vi "无创血糖测量 - OP1.vi"(2 "自动停止(时间, min)":dbl=inf, 3 "自动停止(周期)":dbl=inf, 6 "停止":bool, 8 "每波长测量次数":i32=5) -> ()   [LabVIEW 2026, in "UI-无创.lvlib"]
doc: "演示在LabVIEW中使用队列消息处理器设计模式的基本概念。最简单的队列消息处理器由2个循环组成。“事件处理”循环通过消息队列，将用户界面事件排序为消息队列。这些消息在“消息处理”循环中出队列。注意，“消息处理”循环可以发送消息到自身。"
uses:
  Supports/Sample Settings.ctl
  Supports/Time and Data_OP.ctl
  Supports/Indicators.ctl
  Supports/Save Delay.ctl
  Supports/Wait.ctl
  edcda3f2-1f62-46c4-afbc-dd8e26708560.vi
  <userlib>/_NEVSTOP/Communicable State Machine(CSM)/_Polymophic/CSM - Filter Duplicated Lines.vi
  bab69f4f-9fd6-417e-a657-ac8894b0f8d8.vi
  d5895689-cc80-4a4a-a33c-9882731dfd02.vi
  f416c2de-9cb5-4443-bebf-7c1bee069e61.vi
  fd816077-8d56-410d-a0c7-cc4ae2a0e191.vi
  08ddb0b4-3b06-4116-9f05-deeb9bd3c211.vi
  061f1162-64f0-4531-a8c2-9a7eea5321b3.vi
  09afc524-d839-46af-9592-a0aacb215298.vi
  5ba6a803-8b84-4c90-b72e-7e276277037c.vi
  b6cdf660-3919-45d4-85c6-d3657d11d8bc.vi
  f8a7c933-f379-43a8-9cf8-4111b079c53a.vi
  718ea2b6-ff8b-423b-986a-2c170ecbcd93.vi
  8d110828-7224-455b-9905-edcb614ae088.vi
  4370ed70-8aad-4095-b2cf-34cad3ed2884.vi
  f8ba2474-ccb7-423d-8431-6c03567d15cf.vi
  a0d9968b-1639-45b9-bbc0-305e148ad7f7.vi
  cb0edb06-5019-4007-b477-f13abbf19ffa.vi
  247eb9d3-7548-4bf8-b62b-528284e886c2.vi
  4376c9b7-509c-471f-b1d3-8cb46ece328f.vi
  de3643d5-93ce-4497-bc99-e27b2e615104.vi
  9461128d-940e-41b1-9239-c78715a8a9a5.vi
  <userlib>/_NEVSTOP/Communicable State Machine(CSM)/_Polymophic/CSM - Replace Marks in Messages.vi
  25bd028a-d17a-46b4-b21d-632ed2f3469a.vi
  d2b4f8cd-6edf-4211-ac58-cd3e211821b2.vi
  dd4a060d-1cff-4b6c-a087-6a9eb17f14be.vi
  97590eb0-11f5-446d-9d79-d032973c4d82.vi
  a53f6761-35b4-4fd6-839f-3637c2db1062.vi
  819a418a-78a6-4661-8a04-fceb00ec1904.vi
  a7208fe4-f516-4c66-8ccf-1ba7cd583568.vi
  ec42e1cb-42d0-4315-b7d0-8fa8288cf73a.vi
  44771232-a67e-4ac6-a006-f4ca459dacc0.vi
  029717ad-6970-4481-be37-58bd7465a69d.vi
  97b165be-0bc0-4b14-ad3e-a493e446c08a.vi
  1d48b39c-881e-4765-8858-9798fdcca961.vi
  db2b10a7-c803-446c-8216-4c6a8695a7a0.vi
  eafa804a-60e3-4e10-84cb-3ec5a060bb8b.vi
  4c56b258-92b5-47bd-b87e-17d0926c135c.vi
  6ecd949e-e40b-46d1-b377-4bd26220d93a.vi
  2a6fad02-d7d1-4665-9a59-31a169d33988.vi
  5a7fa7cb-8f9b-466d-8ae0-b9117d618831.vi
  c2926f15-ec64-40b8-95a5-1c7032b582cb.vi
  <userlib>/_NEVSTOP/Communicable State Machine(CSM)/AdvanceAPI/CSM - Revert Arguments-Safe String.vi
  <userlib>/_NEVSTOP/Communicable State Machine(CSM)/_Shared/Trim Single-line Text.vi
  <userlib>/_NEVSTOP/Communicable State Machine(CSM)/AdvanceAPI/CSM - Make String Arguments Safe.vi
  <userlib>/_NEVSTOP/Communicable State Machine(CSM)/AdvanceAPI/CSM - Break Down Multiple States String.vi
  <userlib>/_NEVSTOP/Communicable State Machine(CSM)/AdvanceAPI/CSM - Compact Multiple States.vi
  <userlib>/_NEVSTOP/Communicable State Machine(CSM)/_Shared/Remove Comments from Single-line.vi
  <userlib>/_NEVSTOP/Communicable State Machine(CSM)/_Shared/Split Single-line Message.vi
  4370ed70-8aad-4095-b2cf-34cad3ed2884.vi/99de0c97-112a-4c86-9094-c187659127e1.vi
  <userlib>/_NEVSTOP/Communicable State Machine(CSM)/Utility/Build Error Cluster.vi
  f8ba2474-ccb7-423d-8431-6c03567d15cf.vi/99de0c97-112a-4c86-9094-c187659127e1.vi
  4376c9b7-509c-471f-b1d3-8cb46ece328f.vi/99de0c97-112a-4c86-9094-c187659127e1.vi
  de3643d5-93ce-4497-bc99-e27b2e615104.vi/99de0c97-112a-4c86-9094-c187659127e1.vi
  <userlib>/_NEVSTOP/Communicable State Machine(CSM)/AdvanceAPI/CSM - Keywords.vi
  <userlib>/_NEVSTOP/Communicable State Machine(CSM)/addons/INI-Static-Variable-Support/_Support/instances/_CSM - Read File Logger Configuration - v1.0.vi
  <vilib>/Utility/Data Type/Get Type Information.vi
  <userlib>/_NEVSTOP/Communicable State Machine(CSM)/addons/API-String-Arugments-Support/_Support/Data To SingleElementsArray_csm.vi
  <userlib>/_NEVSTOP/Communicable State Machine(CSM)/addons/API-String-Arugments-Support/_Support/Data To API String Arguments.vi
  <userlib>/_NEVSTOP/Communicable State Machine(CSM)/addons/INI-Static-Variable-Support/_Support/Parse Used Session and Name.vi
  <userlib>/_NEVSTOP/Communicable State Machine(CSM)/addons/INI-Static-Variable-Support/_Support/INI-FGV(lvlibp).vi
  <userlib>/_NEVSTOP/Communicable State Machine(CSM)/addons/INI-Static-Variable-Support/_Support/Populate String with INI Variable.vi
  <userlib>/_NEVSTOP/Communicable State Machine(CSM)/addons/API-String-Arugments-Support/_Support/Convert API String Arguments to Data(variant).vi
  <userlib>/_NEVSTOP/Communicable State Machine(CSM)/addons/API-String-Arugments-Support/_Support/SingleElementsArray To Data_csm.vi
  <userlib>/_NEVSTOP/Communicable State Machine(CSM)/AdvanceAPI/CSM - Get Module Attribute.vi
  <userlib>/_NEVSTOP/Communicable State Machine(CSM)/addons/MassData-Parameter/_support/FGV-MassData(lvlibp).vi
  <userlib>/_NEVSTOP/Communicable State Machine(CSM)/AdvanceAPI/CSM - Set Module Attribute.vi
  <vilib>/express/express arith-compare/Formula/XNode/ExpressFormulaBlockNode.xnode
  <vilib>/Analysis/NI_AALBase.lvlib
  <userlib>/_NEVSTOP/Communicable State Machine(CSM)/Communicable State Machine.lvlib
  Acquisition/Acquisition.lvlib
  Logging/Logging.lvlib
  <userlib>/_NEVSTOP/Communicable State Machine(CSM)/addons/INI-Static-Variable-Support/INI-Static-Variable-Support.lvlib
  <userlib>/_NEVSTOP/Communicable State Machine(CSM)/addons/MassData-Parameter/CSM MassData Parameter Support.lvlib
  <userlib>/_NEVSTOP/Communicable State Machine(CSM)/addons/Watchdog/CSM Watchdog.lvlib
  <userlib>/_NEVSTOP/Communicable State Machine(CSM)/addons/Logger/CSM File Logger.lvlib
  <vilib>/gmath/NI_Gmath.lvlib
panel:
  in  "CSM Name":string="OP1"
  in  "开始":bool
  in  "波形查看":T1(tab)=enum."长期 单环B"
  out "1213":dbl[](graph)
  out "1314":dbl[](graph)
  out "1409":dbl[](graph)
  out "1550":dbl[](graph)
  out "1609":dbl[](graph)
  out "1050":dbl[](graph)
  out "1050 2":dbl[](graph)
  out "1213 3":dbl[](graph)
  out "1314 2":dbl[](graph)
  out "1409 3":dbl[](graph)
  out "1550 3":dbl[](graph)
  out "1609 3":dbl[](graph)
  out "1050":dbl[](graph)=[nan, nan, nan, nan, nan, nan, nan, nan, nan, nan, nan, nan, nan, nan, nan, nan, nan, nan, nan, nan, nan, nan, nan, nan]
  out "1213":dbl[](graph)=[nan, nan, nan, nan, nan, nan, nan, nan, nan, nan, nan, nan, nan, nan, nan, nan, nan, nan, nan, nan, nan, nan, nan, nan]
  out "1314":dbl[](graph)=[nan, nan, nan, nan, nan, nan, nan, nan, nan, nan, nan, nan, nan, nan, nan, nan, nan, nan, nan, nan, nan, nan, nan, nan]
  out "1409":dbl[](graph)=[nan, nan, nan, nan, nan, nan, nan, nan, nan, nan, nan, nan, nan, nan, nan, nan, nan]
  out "1550":dbl[](graph)=[nan, nan, nan, nan, nan, nan, nan, nan, nan, nan, nan, nan]
  out "1609":dbl[](graph)=[nan, nan, nan, nan, nan, nan, nan, nan, nan, nan, nan, nan]
  out "1050 3":dbl[](graph)
  out "1213 2":dbl[](graph)
  out "1314 3":dbl[](graph)
  out "1409 2":dbl[](graph)
  out "1550 2":dbl[](graph)
  out "1609 2":dbl[](graph)
  out "1050 4":dbl[](graph)
  out "1213 4":dbl[](graph)
  out "1314 4":dbl[](graph)
  out "1409 4":dbl[](graph)
  out "1550 4":dbl[](graph)
  out "1609 4":dbl[](graph)
  out "1609 5":dbl[](graph)
  out "1550 5":dbl[](graph)
  out "1409 5":dbl[](graph)
  out "1314 5":dbl[](graph)
  out "1213 5":dbl[](graph)
  out "1050 5":dbl[](graph)
  out "1050 16":dbl[](graph)
  out "1213 16":dbl[](graph)
  out "1314 16":dbl[](graph)
  out "1409 16":dbl[](graph)
  out "1550 14":dbl[](graph)
  out "1609 16":dbl[](graph)
  out "1609 15":dbl[](graph)
  out "1550 9":dbl[](graph)
  out "1409 15":dbl[](graph)
  out "1314 15":dbl[](graph)
  out "1213 15":dbl[](graph)
  out "1050 15":dbl[](graph)
  out "1050 6":dbl[](graph)=[nan, nan, nan, nan, nan, nan, nan, nan, nan, nan, nan, nan, nan, nan, nan, nan, nan, nan, nan, nan, nan, nan, nan, nan]
  out "1213 6":dbl[](graph)=[nan, nan, nan, nan, nan, nan, nan, nan, nan, nan, nan, nan, nan, nan, nan, nan, nan, nan, nan, nan, nan, nan, nan, nan]
  out "1314 6":dbl[](graph)=[nan, nan, nan, nan, nan, nan, nan, nan, nan, nan, nan, nan, nan, nan, nan, nan, nan, nan, nan, nan, nan, nan, nan, nan]
  out "1409 6":dbl[](graph)=[nan, nan, nan, nan, nan, nan, nan, nan, nan, nan, nan, nan, nan, nan, nan, nan, nan]
  out "1550 6":dbl[](graph)=[nan, nan, nan, nan, nan, nan, nan, nan, nan, nan, nan, nan]
  out "1609 6":dbl[](graph)=[nan, nan, nan, nan, nan, nan, nan, nan, nan, nan, nan, nan]
  out "1050 7":dbl[](graph)=[nan, nan, nan, nan, nan, nan, nan, nan, nan, nan, nan, nan, nan, nan, nan, nan, nan, nan, nan, nan, nan, nan, nan, nan]
  out "1213 7":dbl[](graph)=[nan, nan, nan, nan, nan, nan, nan, nan, nan, nan, nan, nan, nan, nan, nan, nan, nan, nan, nan, nan, nan, nan, nan, nan]
  out "1314 7":dbl[](graph)=[nan, nan, nan, nan, nan, nan, nan, nan, nan, nan, nan, nan, nan, nan, nan, nan, nan, nan, nan, nan, nan, nan, nan, nan]
  out "1409 7":dbl[](graph)=[nan, nan, nan, nan, nan, nan, nan, nan, nan, nan, nan, nan, nan, nan, nan, nan, nan]
  out "1550 7":dbl[](graph)=[nan, nan, nan, nan, nan, nan, nan, nan, nan, nan, nan, nan]
  out "1609 7":dbl[](graph)=[nan, nan, nan, nan, nan, nan, nan, nan, nan, nan, nan, nan]
  out "1050 8":dbl[](graph)=[nan, nan, nan, nan, nan, nan, nan, nan, nan, nan, nan, nan, nan, nan, nan, nan, nan, nan, nan, nan, nan, nan, nan, nan]
  out "1213 8":dbl[](graph)=[nan, nan, nan, nan, nan, nan, nan, nan, nan, nan, nan, nan, nan, nan, nan, nan, nan, nan, nan, nan, nan, nan, nan, nan]
  out "1314 8":dbl[](graph)=[nan, nan, nan, nan, nan, nan, nan, nan, nan, nan, nan, nan, nan, nan, nan, nan, nan, nan, nan, nan, nan, nan, nan, nan]
  out "1409 8":dbl[](graph)=[nan, nan, nan, nan, nan, nan, nan, nan, nan, nan, nan, nan, nan, nan, nan, nan, nan]
  out "1550 8":dbl[](graph)=[nan, nan, nan, nan, nan, nan, nan, nan, nan, nan, nan, nan]
  out "1609 8":dbl[](graph)=[nan, nan, nan, nan, nan, nan, nan, nan, nan, nan, nan, nan]
  out "1050 12":dbl[](graph)=[nan, nan, nan, nan, nan, nan, nan, nan, nan, nan, nan, nan, nan, nan, nan, nan, nan, nan, nan, nan, nan, nan, nan, nan]
  out "1213 12":dbl[](graph)=[nan, nan, nan, nan, nan, nan, nan, nan, nan, nan, nan, nan, nan, nan, nan, nan, nan, nan, nan, nan, nan, nan, nan, nan]
  out "1314 12":dbl[](graph)=[nan, nan, nan, nan, nan, nan, nan, nan, nan, nan, nan, nan, nan, nan, nan, nan, nan, nan, nan, nan, nan, nan, nan, nan]
  out "1409 12":dbl[](graph)=[nan, nan, nan, nan, nan, nan, nan, nan, nan, nan, nan, nan, nan, nan, nan, nan, nan]
  out "1550 12":dbl[](graph)=[nan, nan, nan, nan, nan, nan, nan, nan, nan, nan, nan, nan]
  out "1609 12":dbl[](graph)=[nan, nan, nan, nan, nan, nan, nan, nan, nan, nan, nan, nan]
  out "1050 13":dbl[](graph)=[nan, nan, nan, nan, nan, nan, nan, nan, nan, nan, nan, nan, nan, nan, nan, nan, nan, nan, nan, nan, nan, nan, nan, nan]
  out "1213 13":dbl[](graph)=[nan, nan, nan, nan, nan, nan, nan, nan, nan, nan, nan, nan, nan, nan, nan, nan, nan, nan, nan, nan, nan, nan, nan, nan]
  out "1314 13":dbl[](graph)=[nan, nan, nan, nan, nan, nan, nan, nan, nan, nan, nan, nan, nan, nan, nan, nan, nan, nan, nan, nan, nan, nan, nan, nan]
  out "1409 13":dbl[](graph)=[nan, nan, nan, nan, nan, nan, nan, nan, nan, nan, nan, nan, nan, nan, nan, nan, nan]
  out "1550 13":dbl[](graph)=[nan, nan, nan, nan, nan, nan, nan, nan, nan, nan, nan, nan]
  out "1609 13":dbl[](graph)=[nan, nan, nan, nan, nan, nan, nan, nan, nan, nan, nan, nan]
  out "1050 14":dbl[](graph)=[nan, nan, nan, nan, nan, nan, nan, nan, nan, nan, nan, nan, nan, nan, nan, nan, nan, nan, nan, nan, nan, nan, nan, nan]
  out "1213 14":dbl[](graph)=[nan, nan, nan, nan, nan, nan, nan, nan, nan, nan, nan, nan, nan, nan, nan, nan, nan, nan, nan, nan, nan, nan, nan, nan]
  out "1314 14":dbl[](graph)=[nan, nan, nan, nan, nan, nan, nan, nan, nan, nan, nan, nan, nan, nan, nan, nan, nan, nan, nan, nan, nan, nan, nan, nan]
  out "1409 14":dbl[](graph)=[nan, nan, nan, nan, nan, nan, nan, nan, nan, nan, nan, nan, nan, nan, nan, nan, nan]
  out "1550 24":dbl[](graph)=[nan, nan, nan, nan, nan, nan, nan, nan, nan, nan, nan, nan]
  out "1609 14":dbl[](graph)=[nan, nan, nan, nan, nan, nan, nan, nan, nan, nan, nan, nan]
  out "1050 9":dbl[](graph)=[nan, nan, nan, nan, nan, nan, nan, nan, nan, nan, nan, nan, nan, nan, nan, nan, nan, nan, nan, nan, nan, nan, nan, nan]
  out "1213 9":dbl[](graph)=[nan, nan, nan, nan, nan, nan, nan, nan, nan, nan, nan, nan, nan, nan, nan, nan, nan, nan, nan, nan, nan, nan, nan, nan]
  out "1314 9":dbl[](graph)=[nan, nan, nan, nan, nan, nan, nan, nan, nan, nan, nan, nan, nan, nan, nan, nan, nan, nan, nan, nan, nan, nan, nan, nan]
  out "1409 9":dbl[](graph)=[nan, nan, nan, nan, nan, nan, nan, nan, nan, nan, nan, nan, nan, nan, nan, nan, nan]
  out "1550 45":dbl[](graph)=[nan, nan, nan, nan, nan, nan, nan, nan, nan, nan, nan, nan]
  out "1609 9":dbl[](graph)=[nan, nan, nan, nan, nan, nan, nan, nan, nan, nan, nan, nan]
  out "1050 10":dbl[](graph)=[nan, nan, nan, nan, nan, nan, nan, nan, nan, nan, nan, nan, nan, nan, nan, nan, nan, nan, nan, nan, nan, nan, nan, nan]
  out "1213 10":dbl[](graph)=[nan, nan, nan, nan, nan, nan, nan, nan, nan, nan, nan, nan, nan, nan, nan, nan, nan, nan, nan, nan, nan, nan, nan, nan]
  out "1314 10":dbl[](graph)=[nan, nan, nan, nan, nan, nan, nan, nan, nan, nan, nan, nan, nan, nan, nan, nan, nan, nan, nan, nan, nan, nan, nan, nan]
  out "1409 10":dbl[](graph)=[nan, nan, nan, nan, nan, nan, nan, nan, nan, nan, nan, nan, nan, nan, nan, nan, nan]
  out "1550 10":dbl[](graph)=[nan, nan, nan, nan, nan, nan, nan, nan, nan, nan, nan, nan]
  out "1609 10":dbl[](graph)=[nan, nan, nan, nan, nan, nan, nan, nan, nan, nan, nan, nan]
  out "1050 11":dbl[](graph)=[nan, nan, nan, nan, nan, nan, nan, nan, nan, nan, nan, nan, nan, nan, nan, nan, nan, nan, nan, nan, nan, nan, nan, nan]
  out "1213 11":dbl[](graph)=[nan, nan, nan, nan, nan, nan, nan, nan, nan, nan, nan, nan, nan, nan, nan, nan, nan, nan, nan, nan, nan, nan, nan, nan]
  out "1314 11":dbl[](graph)=[nan, nan, nan, nan, nan, nan, nan, nan, nan, nan, nan, nan, nan, nan, nan, nan, nan, nan, nan, nan, nan, nan, nan, nan]
  out "1409 11":dbl[](graph)=[nan, nan, nan, nan, nan, nan, nan, nan, nan, nan, nan, nan, nan, nan, nan, nan, nan]
  out "1550 11":dbl[](graph)=[nan, nan, nan, nan, nan, nan, nan, nan, nan, nan, nan, nan]
  out "1609 11":dbl[](graph)=[nan, nan, nan, nan, nan, nan, nan, nan, nan, nan, nan, nan]
  out "1050 20":dbl[](graph)
  out "1213 20":dbl[](graph)
  out "1314 20":dbl[](graph)
  out "1409 20":dbl[](graph)
  out "1550 18":dbl[](graph)
  out "1609 20":dbl[](graph)
  out "1050 19":dbl[](graph)
  out "1213 19":dbl[](graph)
  out "1314 19":dbl[](graph)
  out "1409 19":dbl[](graph)
  out "1550 17":dbl[](graph)
  out "1609 19":dbl[](graph)
  out "1609 18":dbl[](graph)
  out "1550 16":dbl[](graph)
  out "1409 18":dbl[](graph)
  out "1314 18":dbl[](graph)
  out "1213 18":dbl[](graph)
  out "1050 18":dbl[](graph)
  out "1050 23":dbl[](graph)
  out "1213 23":dbl[](graph)
  out "1314 23":dbl[](graph)
  out "1409 23":dbl[](graph)
  out "1550 21":dbl[](graph)
  out "1609 23":dbl[](graph)
  out "1050 22":dbl[](graph)
  out "1213 22":dbl[](graph)
  out "1314 22":dbl[](graph)
  out "1409 22":dbl[](graph)
  out "1550 20":dbl[](graph)
  out "1609 22":dbl[](graph)
  out "1609 21":dbl[](graph)
  out "1550 19":dbl[](graph)
  out "1409 21":dbl[](graph)
  out "1314 21":dbl[](graph)
  out "1213 21":dbl[](graph)
  out "1050 21":dbl[](graph)
  out "1050 26":dbl[](graph)
  out "1213 26":dbl[](graph)
  out "1314 26":dbl[](graph)
  out "1409 26":dbl[](graph)
  out "1550 25":dbl[](graph)
  out "1609 26":dbl[](graph)
  out "1050 25":dbl[](graph)
  out "1213 25":dbl[](graph)
  out "1314 25":dbl[](graph)
  out "1409 25":dbl[](graph)
  out "1550 23":dbl[](graph)
  out "1609 25":dbl[](graph)
  out "1609 24":dbl[](graph)
  out "1550 22":dbl[](graph)
  out "1409 24":dbl[](graph)
  out "1314 24":dbl[](graph)
  out "1213 24":dbl[](graph)
  out "1050 24":dbl[](graph)
  out "1609 27":dbl[](graph)
  out "1550 26":dbl[](graph)
  out "1409 27":dbl[](graph)
  out "1314 27":dbl[](graph)
  out "1213 27":dbl[](graph)
  out "1050 27":dbl[](graph)
  out "1609 17":dbl[](graph)
  out "1550 15":dbl[](graph)
  out "1409 17":dbl[](graph)
  out "1314 17":dbl[](graph)
  out "1213 17":dbl[](graph)
  out "1050 17":dbl[](graph)
  in  "单环Aa":T2=4 items=["1", "2", "3", "4", "5", "6", "7"]
  out "N单环Ac":dbl
  out "N单环Ab":dbl
  out "N单环Aa":dbl
  out "F单环Ac":dbl[](graph)
  out "F单环Ab":dbl[](graph)
  out "F单环Aa":dbl[][](graph)
  in  "W单环Aa":T3 items=["1050", "1213", "1314", "1409", "1550", "1609"]
  in  "W单环Ab":T3=1 items=["1050", "1213", "1314", "1409", "1550", "1609"]
  in  "W单环Ac":T3=2 items=["1050", "1213", "1314", "1409", "1550", "1609"]
  in  "单环Ac":T2=4 items=["1", "2", "3", "4", "5", "6", "7"]
  in  "单环Ab":T2=4 items=["1", "2", "3", "4", "5", "6", "7"]
  in  "单环Ba":T2=4 items=["1", "2", "3", "4", "5", "6", "7"]
  out "N单环Bc":dbl
  out "N单环Bb":dbl
  out "N单环Ba":dbl
  out "F单环Bc":dbl[](graph)
  out "F单环Bb":dbl[](graph)
  out "F单环Ba":dbl[][](graph)
  in  "W单环Ba":T3=3 items=["1050", "1213", "1314", "1409", "1550", "1609"]
  in  "W单环Bb":T3=4 items=["1050", "1213", "1314", "1409", "1550", "1609"]
  in  "W单环Bc":T3=5 items=["1050", "1213", "1314", "1409", "1550", "1609"]
  in  "单环Bc":T2=4 items=["1", "2", "3", "4", "5", "6", "7"]
  in  "单环Bb":T2=4 items=["1", "2", "3", "4", "5", "6", "7"]
  in  "单环Ca":T2=2 items=["1", "2", "3", "4", "5", "6", "7"]
  out "N单环Cc":dbl
  out "N单环Cb":dbl
  out "N单环Ca":dbl
  out "F单环Cc":dbl[](graph)
  out "F单环Cb":dbl[](graph)
  out "F单环Ca":dbl[][](graph)
  in  "W单环Ca":T3=4 items=["1050", "1213", "1314", "1409", "1550", "1609"]
  in  "W单环Cb":T3=4 items=["1050", "1213", "1314", "1409", "1550", "1609"]
  in  "W单环Cc":T3=4 items=["1050", "1213", "1314", "1409", "1550", "1609"]
  in  "单环Cc":T2=4 items=["1", "2", "3", "4", "5", "6", "7"]
  in  "单环Cb":T2=3 items=["1", "2", "3", "4", "5", "6", "7"]
  in  "R单环Aa":bool
  in  "R单环Ac":bool
  in  "R单环Ab":bool
  in  "R单环Ba":bool
  in  "R单环Bc":bool
  in  "R单环Ca":bool
  in  "R单环Cc":bool
  in  "R单环Bb":bool
  in  "R单环Cb":bool
  in  "R差分Aa":bool
  in  "R差分Ab":bool
  in  "R差分Ac":bool
  in  "R差分Bb":bool
  in  "R差分Bc":bool
  in  "R差分Ba":bool
  in  "R差分Ca":bool
  in  "R差分Cb":bool
  in  "R差分Cc":bool
  in  "R差分Da":bool
  in  "R差分Db":bool
  in  "R差分Dc":bool
  in  "R差分Ea":bool
  in  "R差分Eb":bool
  in  "R差分Ec":bool
  in  "R差分Fa":bool
  in  "R差分Fb":bool
  in  "R差分Fc":bool
  in  "R差分Ga":bool
  in  "R差分Gb":bool
  in  "R差分Gc":bool
  in  "R差分Ha":bool
  in  "R差分Hb":bool
  in  "R差分Hc":bool
  in  "波长差分A":bool
  in  "波长差分B":bool
  in  "波长差分A2":bool
  in  "波长差分B2":bool
  in  "波长差分B3":bool
  in  "波长差分A3":bool
  out "N差分Ac":dbl=nan
  out "N差分Ab":dbl=nan
  out "N差分Aa":dbl=nan
  out "F差分Ac":dbl[](graph)
  out "F差分Ab":dbl[](graph)
  out "F差分Aa":dbl[][](graph)
  in  "W差分Aa":T3 items=["1050", "1213", "1314", "1409", "1550", "1609"]
  in  "W差分Ab":T3 items=["1050", "1213", "1314", "1409", "1550", "1609"]
  in  "W差分Ac":T3 items=["1050", "1213", "1314", "1409", "1550", "1609"]
  in  "差分Aa":T4=9 items=["1-2", "1-3", "1-4", "1-5", "2-3", "2-4", "2-5", "3-4", "3-5", "4-5", "1-6", "1-7", "2-6", "2-7", "3-6", "3-7", "4-6", "4-7", "5-6", "5-7", "6-7"]
  in  "差分Ab":T4=7 items=["1-2", "1-3", "1-4", "1-5", "2-3", "2-4", "2-5", "3-4", "3-5", "4-5", "1-6", "1-7", "2-6", "2-7", "3-6", "3-7", "4-6", "4-7", "5-6", "5-7", "6-7"]
  in  "差分Ac":T4=4 items=["1-2", "1-3", "1-4", "1-5", "2-3", "2-4", "2-5", "3-4", "3-5", "4-5", "1-6", "1-7", "2-6", "2-7", "3-6", "3-7", "4-6", "4-7", "5-6", "5-7", "6-7"]
  out "N差分Bc":dbl=nan
  out "N差分Bb":dbl=nan
  out "N差分Ba":dbl=nan
  out "F差分Bc":dbl[](graph)
  out "F差分Bb":dbl[](graph)
  out "F差分Ba":dbl[][](graph)
  in  "W差分Ba":T3=1 items=["1050", "1213", "1314", "1409", "1550", "1609"]
  in  "W差分Bb":T3=1 items=["1050", "1213", "1314", "1409", "1550", "1609"]
  in  "W差分Bc":T3=1 items=["1050", "1213", "1314", "1409", "1550", "1609"]
  in  "差分Bc":T4=4 items=["1-2", "1-3", "1-4", "1-5", "2-3", "2-4", "2-5", "3-4", "3-5", "4-5", "1-6", "1-7", "2-6", "2-7", "3-6", "3-7", "4-6", "4-7", "5-6", "5-7", "6-7"]
  in  "差分Bb":T4=7 items=["1-2", "1-3", "1-4", "1-5", "2-3", "2-4", "2-5", "3-4", "3-5", "4-5", "1-6", "1-7", "2-6", "2-7", "3-6", "3-7", "4-6", "4-7", "5-6", "5-7", "6-7"]
  in  "差分Ba":T4=9 items=["1-2", "1-3", "1-4", "1-5", "2-3", "2-4", "2-5", "3-4", "3-5", "4-5", "1-6", "1-7", "2-6", "2-7", "3-6", "3-7", "4-6", "4-7", "5-6", "5-7", "6-7"]
  out "N差分Cc":dbl=nan
  out "N差分Cb":dbl=nan
  out "N差分Ca":dbl=nan
  out "F差分Cc":dbl[](graph)
  out "F差分Cb":dbl[](graph)
  out "F差分Ca":dbl[][](graph)
  in  "W差分Ca":T3=2 items=["1050", "1213", "1314", "1409", "1550", "1609"]
  in  "W差分Cb":T3=2 items=["1050", "1213", "1314", "1409", "1550", "1609"]
  in  "W差分Cc":T3=2 items=["1050", "1213", "1314", "1409", "1550", "1609"]
  in  "差分Cc":T4=4 items=["1-2", "1-3", "1-4", "1-5", "2-3", "2-4", "2-5", "3-4", "3-5", "4-5", "1-6", "1-7", "2-6", "2-7", "3-6", "3-7", "4-6", "4-7", "5-6", "5-7", "6-7"]
  in  "差分Ca":T4=9 items=["1-2", "1-3", "1-4", "1-5", "2-3", "2-4", "2-5", "3-4", "3-5", "4-5", "1-6", "1-7", "2-6", "2-7", "3-6", "3-7", "4-6", "4-7", "5-6", "5-7", "6-7"]
  in  "差分Cb":T4=7 items=["1-2", "1-3", "1-4", "1-5", "2-3", "2-4", "2-5", "3-4", "3-5", "4-5", "1-6", "1-7", "2-6", "2-7", "3-6", "3-7", "4-6", "4-7", "5-6", "5-7", "6-7"]
  out "N差分Dc":dbl=nan
  out "N差分Db":dbl=nan
  out "N差分Da":dbl=nan
  out "F差分Dc":dbl[](graph)
  out "F差分Db":dbl[](graph)
  out "F差分Da":dbl[][](graph)
  in  "W差分Da":T3=3 items=["1050", "1213", "1314", "1409", "1550", "1609"]
  in  "W差分Db":T3=3 items=["1050", "1213", "1314", "1409", "1550", "1609"]
  in  "W差分Dc":T3=3 items=["1050", "1213", "1314", "1409", "1550", "1609"]
  in  "差分Da":T4=9 items=["1-2", "1-3", "1-4", "1-5", "2-3", "2-4", "2-5", "3-4", "3-5", "4-5", "1-6", "1-7", "2-6", "2-7", "3-6", "3-7", "4-6", "4-7", "5-6", "5-7", "6-7"]
  in  "差分Db":T4=7 items=["1-2", "1-3", "1-4", "1-5", "2-3", "2-4", "2-5", "3-4", "3-5", "4-5", "1-6", "1-7", "2-6", "2-7", "3-6", "3-7", "4-6", "4-7", "5-6", "5-7", "6-7"]
  in  "差分Dc":T4=4 items=["1-2", "1-3", "1-4", "1-5", "2-3", "2-4", "2-5", "3-4", "3-5", "4-5", "1-6", "1-7", "2-6", "2-7", "3-6", "3-7", "4-6", "4-7", "5-6", "5-7", "6-7"]
  out "N差分Ec":dbl=nan
  out "N差分Eb":dbl=nan
  out "N差分Ea":dbl=nan
  out "F差分Ec":dbl[](graph)
  out "F差分Eb":dbl[](graph)
  out "F差分Ea":dbl[][](graph)
  in  "W差分Ea":T3=4 items=["1050", "1213", "1314", "1409", "1550", "1609"]
  in  "W差分Eb":T3=4 items=["1050", "1213", "1314", "1409", "1550", "1609"]
  in  "W差分Ec":T3=4 items=["1050", "1213", "1314", "1409", "1550", "1609"]
  in  "差分Ea":T4=9 items=["1-2", "1-3", "1-4", "1-5", "2-3", "2-4", "2-5", "3-4", "3-5", "4-5", "1-6", "1-7", "2-6", "2-7", "3-6", "3-7", "4-6", "4-7", "5-6", "5-7", "6-7"]
  in  "差分Eb":T4=7 items=["1-2", "1-3", "1-4", "1-5", "2-3", "2-4", "2-5", "3-4", "3-5", "4-5", "1-6", "1-7", "2-6", "2-7", "3-6", "3-7", "4-6", "4-7", "5-6", "5-7", "6-7"]
  in  "差分Ec":T4=4 items=["1-2", "1-3", "1-4", "1-5", "2-3", "2-4", "2-5", "3-4", "3-5", "4-5", "1-6", "1-7", "2-6", "2-7", "3-6", "3-7", "4-6", "4-7", "5-6", "5-7", "6-7"]
  out "N差分Fc":dbl=nan
  out "N差分Fb":dbl=nan
  out "N差分Fa":dbl=nan
  out "F差分Fc":dbl[](graph)
  out "F差分Fb":dbl[](graph)
  out "F差分Fa":dbl[][](graph)
  in  "W差分Fa":T3=5 items=["1050", "1213", "1314", "1409", "1550", "1609"]
  in  "W差分Fb":T3=5 items=["1050", "1213", "1314", "1409", "1550", "1609"]
  in  "W差分Fc":T3=5 items=["1050", "1213", "1314", "1409", "1550", "1609"]
  in  "差分Fa":T4=9 items=["1-2", "1-3", "1-4", "1-5", "2-3", "2-4", "2-5", "3-4", "3-5", "4-5", "1-6", "1-7", "2-6", "2-7", "3-6", "3-7", "4-6", "4-7", "5-6", "5-7", "6-7"]
  in  "差分Fb":T4=7 items=["1-2", "1-3", "1-4", "1-5", "2-3", "2-4", "2-5", "3-4", "3-5", "4-5", "1-6", "1-7", "2-6", "2-7", "3-6", "3-7", "4-6", "4-7", "5-6", "5-7", "6-7"]
  in  "差分Fc":T4=4 items=["1-2", "1-3", "1-4", "1-5", "2-3", "2-4", "2-5", "3-4", "3-5", "4-5", "1-6", "1-7", "2-6", "2-7", "3-6", "3-7", "4-6", "4-7", "5-6", "5-7", "6-7"]
  out "N差分Gc":dbl=nan
  out "N差分Gb":dbl=nan
  out "N差分Ga":dbl=nan
  out "F差分Gc":dbl[](graph)
  out "F差分Gb":dbl[](graph)
  out "F差分Ga":dbl[][](graph)
  in  "W差分Ga":T3 items=["1050", "1213", "1314", "1409", "1550", "1609"]
  in  "W差分Gb":T3=1 items=["1050", "1213", "1314", "1409", "1550", "1609"]
  in  "W差分Gc":T3=2 items=["1050", "1213", "1314", "1409", "1550", "1609"]
  in  "差分Ga":T4 items=["1-2", "1-3", "1-4", "1-5", "2-3", "2-4", "2-5", "3-4", "3-5", "4-5", "1-6", "1-7", "2-6", "2-7", "3-6", "3-7", "4-6", "4-7", "5-6", "5-7", "6-7"]
  in  "差分Gb":T4 items=["1-2", "1-3", "1-4", "1-5", "2-3", "2-4", "2-5", "3-4", "3-5", "4-5", "1-6", "1-7", "2-6", "2-7", "3-6", "3-7", "4-6", "4-7", "5-6", "5-7", "6-7"]
  in  "差分Gc":T4 items=["1-2", "1-3", "1-4", "1-5", "2-3", "2-4", "2-5", "3-4", "3-5", "4-5", "1-6", "1-7", "2-6", "2-7", "3-6", "3-7", "4-6", "4-7", "5-6", "5-7", "6-7"]
  out "N差分Hc":dbl=nan
  out "N差分Hb":dbl=nan
  out "N差分Ha":dbl=nan
  out "F差分Hc":dbl[](graph)
  out "F差分Hb":dbl[](graph)
  out "F差分Ha":dbl[][](graph)
  in  "W差分Ha":T3=3 items=["1050", "1213", "1314", "1409", "1550", "1609"]
  in  "W差分Hb":T3=4 items=["1050", "1213", "1314", "1409", "1550", "1609"]
  in  "W差分Hc":T3=5 items=["1050", "1213", "1314", "1409", "1550", "1609"]
  in  "差分Ha":T4 items=["1-2", "1-3", "1-4", "1-5", "2-3", "2-4", "2-5", "3-4", "3-5", "4-5", "1-6", "1-7", "2-6", "2-7", "3-6", "3-7", "4-6", "4-7", "5-6", "5-7", "6-7"]
  in  "差分Hb":T4 items=["1-2", "1-3", "1-4", "1-5", "2-3", "2-4", "2-5", "3-4", "3-5", "4-5", "1-6", "1-7", "2-6", "2-7", "3-6", "3-7", "4-6", "4-7", "5-6", "5-7", "6-7"]
  in  "差分Hc":T4 items=["1-2", "1-3", "1-4", "1-5", "2-3", "2-4", "2-5", "3-4", "3-5", "4-5", "1-6", "1-7", "2-6", "2-7", "3-6", "3-7", "4-6", "4-7", "5-6", "5-7", "6-7"]
  in  "k3":dbl=1.0
  in  "差分Y3":T4=8 items=["1-2", "1-3", "1-4", "1-5", "2-3", "2-4", "2-5", "3-4", "3-5", "4-5", "1-6", "1-7", "2-6", "2-7", "3-6", "3-7", "4-6", "4-7", "5-6", "5-7", "6-7"]
  in  "Y3":T3 items=["1050", "1213", "1314", "1409", "1550", "1609"]
  in  "X3":T3=4 items=["1050", "1213", "1314", "1409", "1550", "1609"]
  in  "差分X3":T4=8 items=["1-2", "1-3", "1-4", "1-5", "2-3", "2-4", "2-5", "3-4", "3-5", "4-5", "1-6", "1-7", "2-6", "2-7", "3-6", "3-7", "4-6", "4-7", "5-6", "5-7", "6-7"]
  out "F_dAd_3":dbl[][](graph)
  in  "k2":dbl=1.0
  in  "k":dbl=1.0
  in  "差分Y2":T4=7 items=["1-2", "1-3", "1-4", "1-5", "2-3", "2-4", "2-5", "3-4", "3-5", "4-5", "1-6", "1-7", "2-6", "2-7", "3-6", "3-7", "4-6", "4-7", "5-6", "5-7", "6-7"]
  in  "Y2":T3 items=["1050", "1213", "1314", "1409", "1550", "1609"]
  in  "X2":T3=4 items=["1050", "1213", "1314", "1409", "1550", "1609"]
  in  "差分X2":T4=7 items=["1-2", "1-3", "1-4", "1-5", "2-3", "2-4", "2-5", "3-4", "3-5", "4-5", "1-6", "1-7", "2-6", "2-7", "3-6", "3-7", "4-6", "4-7", "5-6", "5-7", "6-7"]
  in  "差分Y":T4=9 items=["1-2", "1-3", "1-4", "1-5", "2-3", "2-4", "2-5", "3-4", "3-5", "4-5", "1-6", "1-7", "2-6", "2-7", "3-6", "3-7", "4-6", "4-7", "5-6", "5-7", "6-7"]
  out "F_dAd_2":dbl[][](graph)
  out "F_dAd_1":dbl[][](graph)
  in  "Y":T3 items=["1050", "1213", "1314", "1409", "1550", "1609"]
  in  "X":T3=4 items=["1050", "1213", "1314", "1409", "1550", "1609"]
  in  "差分X":T4=9 items=["1-2", "1-3", "1-4", "1-5", "2-3", "2-4", "2-5", "3-4", "3-5", "4-5", "1-6", "1-7", "2-6", "2-7", "3-6", "3-7", "4-6", "4-7", "5-6", "5-7", "6-7"]
  in  "暗电流赋0":bool
  in  "校准模式":T5=enum."逐周期"
  in  "温度校准值（每度）":dbl[][](array[numeric])=[[0.0, 0.0, 0.0, 0.0, 0.0, 0.0, 0.00013, 0.00013, 0.00013, 0.00013, 0.00013, 0.00013], [0.0, 0.0, 0.0, 0.0, 0.0, 0.0, 0.00013, 0.00013, 0.00013, 0.00013, 0.00013, 0.00013], [0.0, 0.0, 0.0, 0.0, 0.0, 0.0, 0.00013, 0.00013, 0.00013, 0.00013, 0.00013, 0.00013], [0.0, 0.0, 0.0, 0.0, 0.0, 0.0, 0.00013, 0.00013, 0.00013, 0.00013, 0.00013, 0.00013], [0.0, 0.0, 0.0, 0.0, 0.0, 0.0, 0.00013, 0.00013, 0.00013, 0.00013, 0.00013, 0.00013], [0.0, 0.0, 0.0, 0.0, 0.0, 0.0, 0.00013, 0.00013, 0.00013, 0.00013, 0.00013, 0.00013], [0.0, 0.0, 0.0, 0.0, 0.0, 0.0, 0.00013, 0.00013, 0.00013, 0.00013, 0.00013, 0.00013], [0.0, 0.0, 0.0, 0.0, 0.0, 0.0, 0.00013, 0.00013, 0.00013, 0.00013, 0.00013, 0.00013], [0.0, 0.0, 0.0, 0.0, 0.0, 0.0, 0.00013, 0.00013, 0.00013, 0.00013, 0.00013, 0.00013], [0.0, 0.0, 0.0, 0.0, 0.0, 0.0, 0.00013, 0.00013, 0.00013, 0.00013, 0.00013, 0.00013], [0.00013, 0.00013, 0.00013, 0.00013, 0.00013, 0.00013, 0.00013, 0.00013, 0.00013, 0.00013, 0.00013, 0.00013], [0.00013, 0.00013, 0.00013, 0.00013, 0.00013, 0.00013, 0.00013, 0.00013, 0.00013, 0.00013, 0.00013, 0.00013], [0.00013, 0.00013, 0.00013, 0.00013, 0.00013, 0.00013, 0.00013, 0.00013, 0.00013, 0.00013, 0.00013, 0.00013], [0.00013, 0.00013, 0.00013, 0.00013, 0.00013, 0.00013, 0.00013, 0.00013, 0.00013, 0.00013, 0.00013, 0.00013], [0.00013, 0.00013, 0.00013, 0.00013, 0.00013, 0.00013, 0.00013, 0.00013, 0.00013, 0.00013, 0.00013, 0.00013], [0.00013, 0.00013, 0.00013, 0.00013, 0.00013, 0.00013, 0.00013, 0.00013, 0.00013, 0.00013, 0.00013, 0.00013], [0.00013, 0.00013, 0.00013, 0.00013, 0.00013, 0.00013, 0.00013, 0.00013, 0.00013, 0.00013, 0.00013, 0.00013], [0.00013, 0.00013, 0.00013, 0.00013, 0.00013, 0.00013, 0.00013, 0.00013, 0.00013, 0.00013, 0.00013, 0.00013], [0.00013, 0.00013, 0.00013, 0.00013, 0.00013, 0.00013, 0.00013, 0.00013, 0.00013, 0.00013, 0.00013, 0.00013], [0.00013, 0.00013, 0.00013, 0.00013, 0.00013, 0.00013, 0.00013, 0.00013, 0.00013, 0.00013, 0.00013, 0.00013]]
  in  "是否校准？":bool
  in  "基准温度":dbl=25.0
  in  "暗电流校准值":dbl[](array[numeric])
  out "校准温度":dbl
  in  "校准通道":T6=enum."温度通道2"
  in  "温度校准系数赋0":bool
  in  "删除项(按曲线编号)":i32
  in  "删除":bool
  out "添加/删除状态":string
  in  "添加":bool
  in  "显示数目":i32=10
  out "45AD":dbl[][](graph)
  out "时间-周期":waveform(i32)(graph)
  out "时间-周期对照":string[][](table) caption="表格"
  out "Error Occurred":errorcluster caption="温度采集-错误输出"
  out "State History":string
  in  "子程序？":bool
  out "State History - Time":string
  in  "测头供电":bool=TRUE
  in  "控制台":enum32{"配置", "控制台", "测量结果", "结果-67环"}(tab)
  in  "光控设备":tag="Dev1"
  in  "测量波长":T3[](array[typedef]) items=["1050", "1213", "1314", "1409", "1550", "1609"]
  in  "等待时":enum16{"无电无光", "有电无光", "无电有光", "有电有光"}(ring)
  in  "等待时间(s)":dbl
  in  "测头类型":T7
  in  "信号采集设备和供电":tag="Dev1"
  in  "数据文件前缀":string
  in  "图表重置":bool
  in  "等待方式":bool
  in  "每x周期/点等待":i32=8 min=0
  in  "计时方式":bool
  in  "测头出光":bool=TRUE
  in  "是否保存":bool
  out "数据保存中？":bool
  in  "差分下限":dbl=-0.002 step=0.001
  in  "差分上限":dbl=0.002 step=0.001
  in  "单环下限":dbl=-0.02 step=0.01
  in  "单环上限":dbl=0.02 step=0.01
  in  "差分图范围":enum32{"自动", "固定", "自定义"}(radio)
  in  "单环图范围":enum32{"自动", "固定", "自定义"}(radio)
  in  "分段颜色":enum32{"蓝色", "红色"}(radio)
  out "计时":string="00: 00: 00"
  in  "暂停/继续":bool=TRUE
  in  "开始/清零":bool
  in  "测头拿取":bool
  out "时间":string="00: 00: 00"
  in  "A | Ad\n基准周期":i32=1
  in  "基准周期设定":bool
  in  "暂停按钮":bool
  in  "重新开始(不改变文件)":bool
  out "已运行时间(min)":dbl=inf format="%.2g"
  out "等待倒计时(s)":dbl format="%.1g"
  out "测量点数(图表)":i32
  out "测量周期":i32
  out "7环SNR":dbl caption="7环"
  out "6环SNR":dbl caption="6环"
  out "7环":dbl format="%0.6f"
  out "6环":dbl format="%0.6f"
  out "2-5":dbl=nan
  out "2-4":dbl=nan
  out "2-3":dbl=nan
  out "1环SNR":dbl caption="1环"
  out "2环SNR":dbl caption="2环"
  out "3环SNR":dbl caption="3环"
  out "4环SNR":dbl caption="4环"
  out "1环":dbl format="%0.6f"
  out "当前周期":i32
  out "当前波长":dbl
  out "第N次测量":i32
  out "2环":dbl format="%0.6f"
  out "3环":dbl format="%0.6f"
  out "4环":dbl format="%0.6f"
  out "波长":i32
  out "1-2":dbl=nan
  out "1-3":dbl=nan
  out "1-4":dbl=nan
  out "5环":dbl format="%0.6f"
  out "5环SNR":dbl caption="5环"
  out "1-5":dbl=nan
  out "3-4":dbl=nan
  out "3-5":dbl=nan
  out "4-5":dbl=nan
  out "6-7":dbl=nan
  out "4-6":dbl=nan
  out "3-7":dbl=nan
  out "3-6":dbl=nan
  out "1-6":dbl=nan
  out "1-7":dbl=nan
  out "2-6":dbl=nan
  out "2-7":dbl=nan
  out "4-7":dbl=nan
  out "5-6":dbl=nan
  out "5-7":dbl=nan
  out "程序状态":string="已停止"
  # "人体无创血糖检测系统---"
  # "1"
  # "2"
  # "1-2"
  # "3"
  # "4"
  # "5"
  # "6"
  # "7"
  # "1-3"
  # "1-4"
  # "1-5"
  # "2-4"
  # "3-5"
  # "2-5"
  # "2-3"
  # "3-4"
  # "4-5"
  # "1-6"
  # "1-7"
  # "2-6"
  # "2-7"
  # "3-6"
  # "3-7"
  # "4-6"
  # "4-7"
  # "5-6"
  # "5-7"
  # "6-7"
  # "X - k*Y"
  # "X - k*Y"
  # "X - k*Y"
  # "1050"
  # "1213"
  # "1314"
  # "1409"
  # "1550"
  # "1609"
  # "5环"
  # "7环"
  # "1-2"
  # "1-2"
  # "1-3"
  # "1-3"
  # "1-4"
  # "1-4"
  # "1环"
  # "1-5"
  # "1-5"
  # "2环"
  # "2-3"
  # "1-6"
  # "3环"
  # "2-4"
  # "1-7"
  # "4环"
  # "2-5"
  # "2-6"
  # "5环"
  # "3-4"
  # "2-7"
  # "6环"
  # "3-5"
  # "3-6"
  # "7环"
  # "4-5"
  # "3-7"
  # "4-6"
  # "4-7"
  # "5-6"
  # "5-7"
  # "6-7"
  # "1050"
  # "1219"
  # "1314"
  # "1409"
  # "1550"
  # "1609"
  # "波长和测量配置"
  # "信号采集和供电"
  # "计时"
  # "添加至旧文件"
  # "(显示和保存)"
  # "时间"
  # "分段颜色"
  # "程序控制"
  # "保存与设备控制"
  # "当前运行信息"
  # "差分"
  # "当前测量数据"
  # "SNR"
  # "单环"
  # "SNR"
  # "差分"
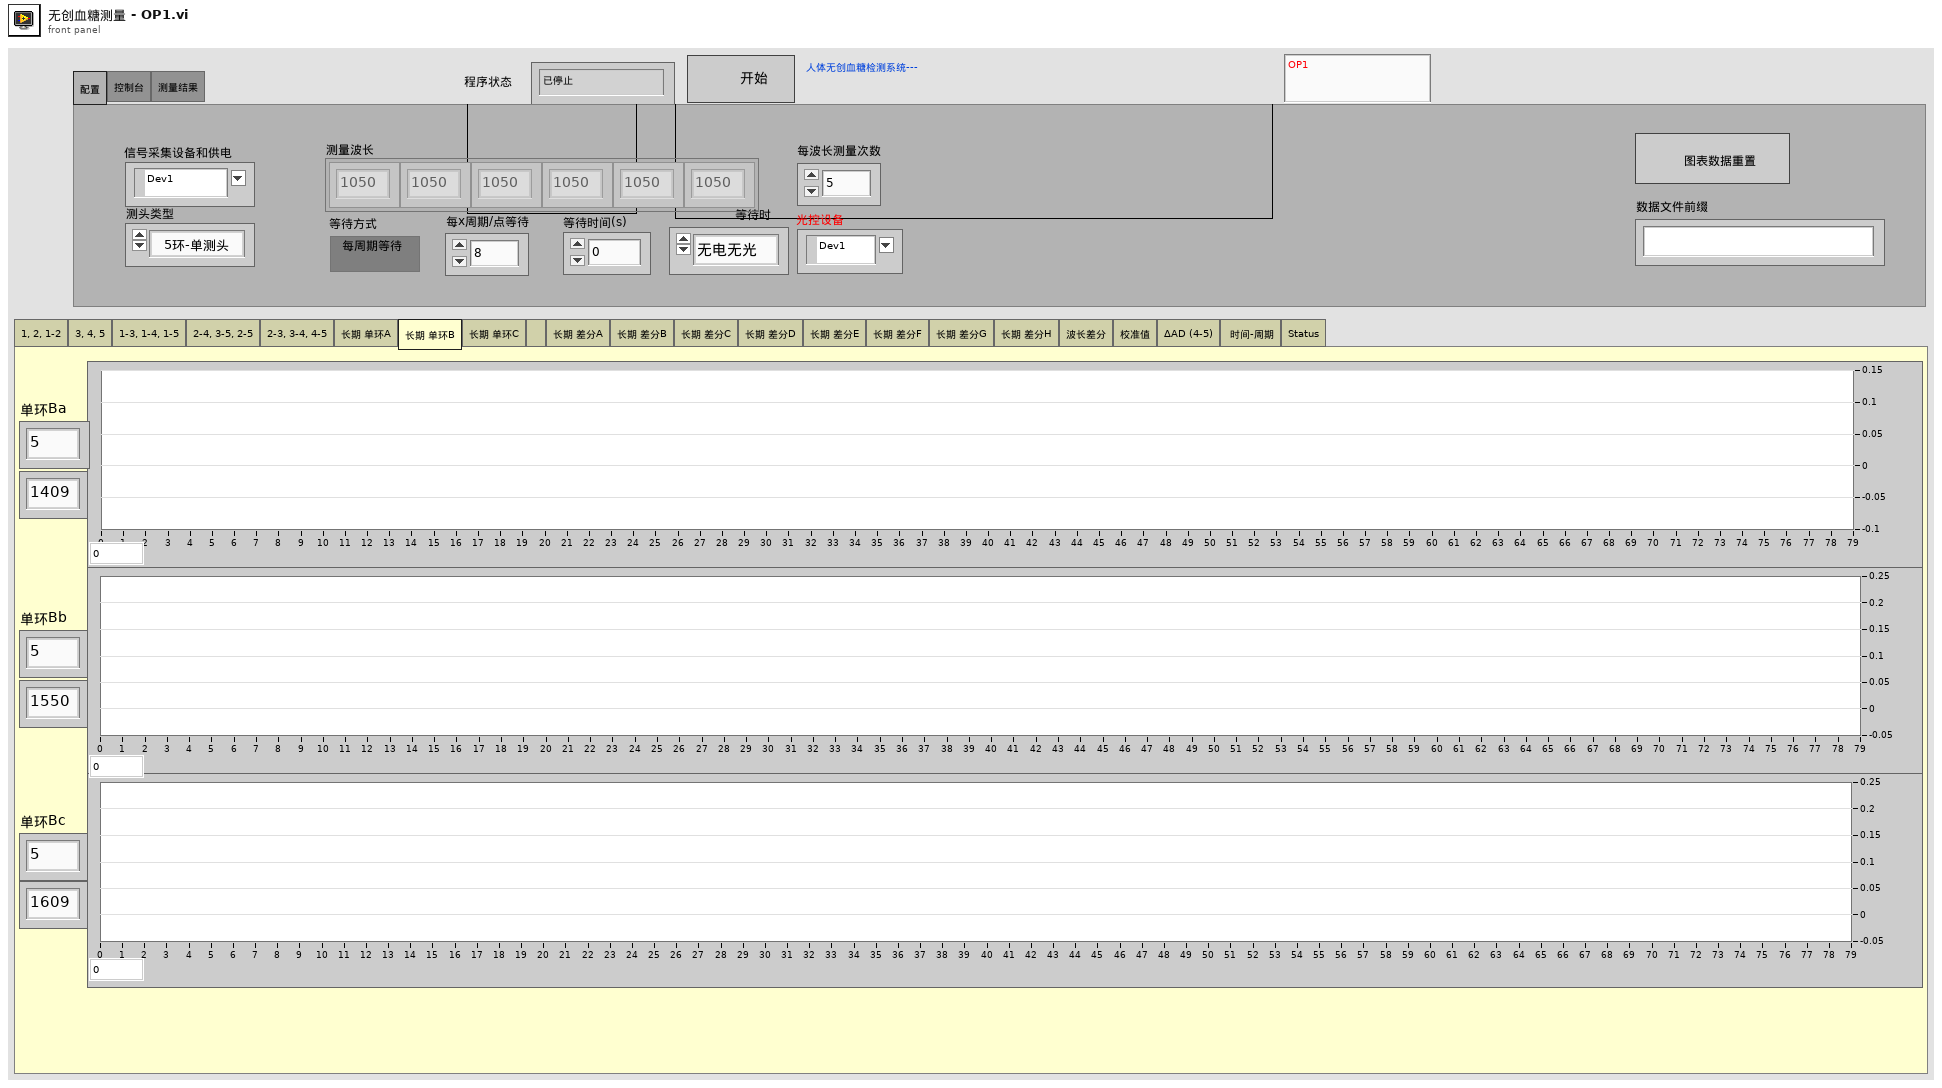
[diagram p1: front panel]
types:
  T1 = enum32{"1, 2, 1-2", "3, 4, 5", "6, 7", "1-3, 1-4, 1-5", "2-4, 3-5, 2-5", "2-3, 3-4, 4-5", "1-6, 1-7, 2-6", "2-7, 3-6, 3-7", "4-6, 4-7, 5-6", "5-7, 6-7", "长期 单环A", "长期 单环B", "长期 单环C", "  ", "长期 差分A", "长期 差分B", "长期 差分C", "长期 差分D", "长期 差分E", "长期 差分F", "长期 差分G", "长期 差分H", "波长差分", "校准值", "ΔAD (4-5)", " 时间-周期", "Status"}
  T2 = typedef "UI-无创.lvlib/单环列表.ctl" = i32
  T3 = typedef "UI-无创.lvlib/波长列表.ctl" = i32
  T4 = typedef "UI-无创.lvlib/差分列表.ctl" = i32
  T5 = typedef "UI-无创.lvlib/暗电流校准模式.ctl" = enum32{"手动", "逐周期"}
  T6 = typedef "温度通道索引_全局.ctl" = enum16{"温度通道1", "温度通道2", "温度通道3", "温度通道4", "温度通道5", "温度通道6", "温度通道7", "温度通道8", "TC1控制温度", "TC1实际温度", "TC1实际输出电压", "TC1实际输出电流", "TC1实际输出功率", "TC2控制温度", "TC2实际温度", "TC2实际输出电压", "TC2实际输出电流", "TC2实际输出功率", "压力(电压值)", "压力(g)", "Zolix当前位置", "Zolix速度", "步进电机位置", "步进电机速度", "温度", "湿度"}
  T7 = typedef "UI-无创.lvlib/测头类型.ctl" = enum16{"5环-单测头", "5环-双测头", "5环-三测头", "7环-单测头", "7环-双测头"}
  T8 = cluster{"Enable":bool, "Limit":cluster{"FileSize":i64, "FileNum":i32}, "Timestamp.Format":string, "AutoExit":bool}
  T9 = enum32{"Invalid", "Standard", "Closed", "Hidden", "Minimized", "Maximized"}
  T10 = enum32{"invalid app kind", "Development System", "Run Time System", "Student Edition", "Embedded LabVIEW", "Evaluation", "Custom"}
  T11 = enum8{"Enabled", "Disabled", "Disabled and Grayed Out"}
  T12 = typedef "UI-无创.lvlib/图表范围自定义.ctl" = cluster{"上限":dbl, "下限":dbl, "图范围":enum32{"自动", "固定", "自定义"}}
  T13 = typedef "UI-无创.lvlib/Save Delay.ctl" = enum16{"Idle", "拿起", "放下-出光", "放下-显示", "放下-保存"}
  T14 = typedef "UI-无创.lvlib/Wait.ctl" = cluster{"每x周期/点等待":i32, "等待方式":bool, "等待时间(s)":dbl, "等待时":enum16{"无电无光", "有电无光", "无电有光", "有电有光"}}
  T15 = typedef "Communicable State Machine.lvlib/_CSM_Response Source Message.ctl" = cluster{"‘State":string, "’Arguments":string, "’Error":errorcluster}
  T16 = cluster{"Current VI Reference":refnum<vi>, "Close Panel on Exit?":bool}
  T17 = typedef "UI-无创.lvlib/Sample Settings.ctl" = cluster{"设备信息":cluster{"初始索引子集":i8[], "模拟信号采集通道":string, "数字-供电":refnum<k21>, "数字-光控":refnum<k21>, "光控设备":tag, "光电设备分离？":bool, "光谱保存路径":path, "环数":u8}, "测量控制":cluster{"测头拿起":bool, "起始保存":bool, "测头供电":bool, "测头出光":bool}, "测量":cluster{"每波长测量次数":i32, "波长":i32[], "起始周期":i32, "起始测量周期":i32}, "等待":cluster{"等待时间(s)":dbl, "等待方式":bool, "每x周期/点等待":i32, "等待时":enum16{"无电无光", "有电无光", "无电有光", "有电有光"}}, "校准":cluster{"暗电流校准值初值":dbl[], "温度校准值":dbl[], "校准模式":T5}, "图表相关":cluster{"文件-时间":string}, "CSM":cluster{"CSM Name":string}}
  T18 = typedef "UI-无创.lvlib/Time and Data_OP.ctl" = cluster{"采集时间":timestamp, "采集时间(dbl)":dbl, "Data":dbl[], "当前运行信息":cluster{"当前周期":i32, "当前次数":i32, "测量周期":i32, "当前索引子集":i8[], "当前波长":i32}, "暗电流校准值":dbl[], "Logging Settings":cluster{"是否保存？":bool, "波长结束？":bool, "周期结束？":bool}, "原始值":cluster{"1环(原始值)":dbl[][], "2环(原始值)":dbl[][], "3环(原始值)":dbl[][], "4环(原始值)":dbl[][], "5环(原始值)":dbl[][], "6环(原始值)":dbl[][], "7环(原始值)":dbl[][]}, "校准值":cluster{"1环(校准值)":dbl[][], "2环(校准值)":dbl[][], "3环(校准值)":dbl[][], "4环(校准值)":dbl[][], "5环(校准值)":dbl[][], "6环(校准值)":dbl[][], "7环(校准值)":dbl[][]}}
  T19 = typedef "UI-无创.lvlib/Indicators.ctl" = cluster{"控制":cluster{"信号采集设备和供电":tag, "自动停止(周期)":dbl, "自动停止(时间, min)":dbl, "测头类型":T7, "测量波长":T3[]}, "校准":cluster{"温度校准值（每度）":dbl[][], "温度校准通道":T6}, "图表相关":cluster{"分段颜色":enum32{"蓝色", "红色"}, "程序开始时间":timestamp, "基准索引":i32}, "Save Delay":cluster{"放下周期":i32, "进度":T13}, "波长差分":cluster{"X":T3, "Y":T3, "差分X":T4, "差分Y":T4, "k":dbl, "X2":T3, "Y2":T3, "差分X2":T4, "差分Y2":T4, "k2":dbl, "X3":T3, "Y3":T3, "差分X3":T4, "差分Y3":T4, "k3":dbl}}
  T20 = cluster{"Core":cluster{"Current VI Reference":refnum<vi>, "Close Panel on Exit?":bool}, "Sample Settings":T17, "Time and Data":T18, "Indicators":T19, "子程序？":bool}
  T21 = typedef "全局变量数据.ctl" = cluster{"温度采集":dbl[], "温度控制":dbl[], "压力测量":dbl[], "Zolix":dbl[], "步进电机":dbl[], "湿度测量":dbl[], "距离测量":dbl[]}
  T22 = cluster{"每x周期/点等待":i32, "等待方式":bool, "等待时间(s)":dbl, "等待时":enum16{"无电无光", "有电无光", "无电有光", "有电有光"}}
  T23 = cluster{"Core":cluster{"Current VI Reference":refnum<vi>, "Close Panel on Exit?":bool}, "Your Boolean data":bool, "Your string data":string}
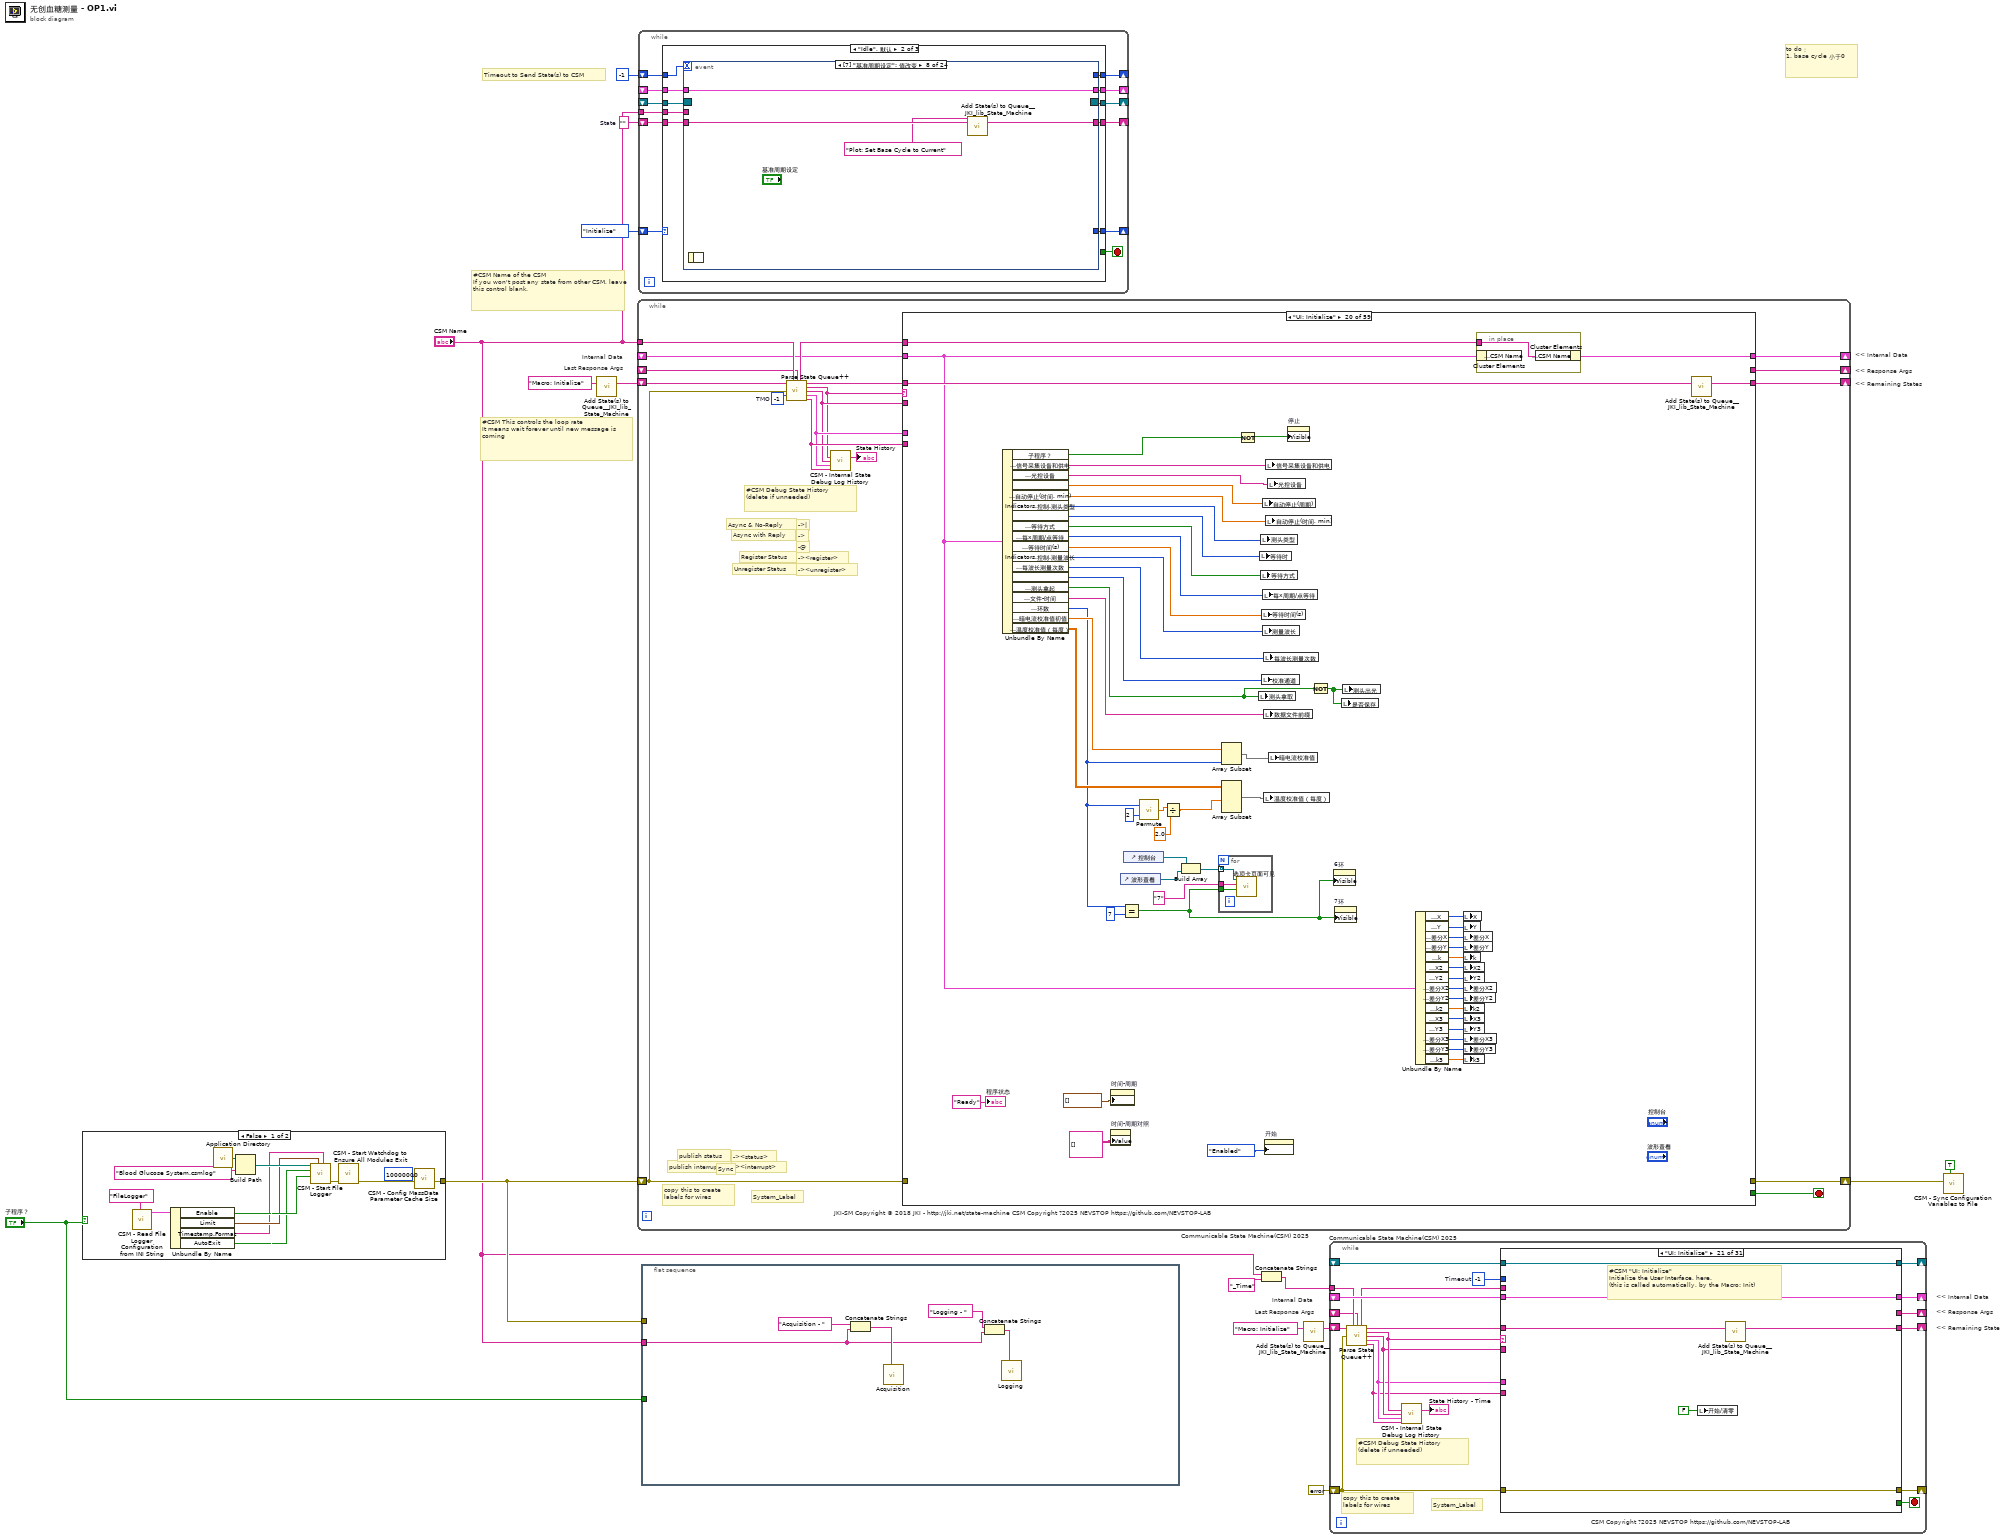
[diagram p0: block diagram]
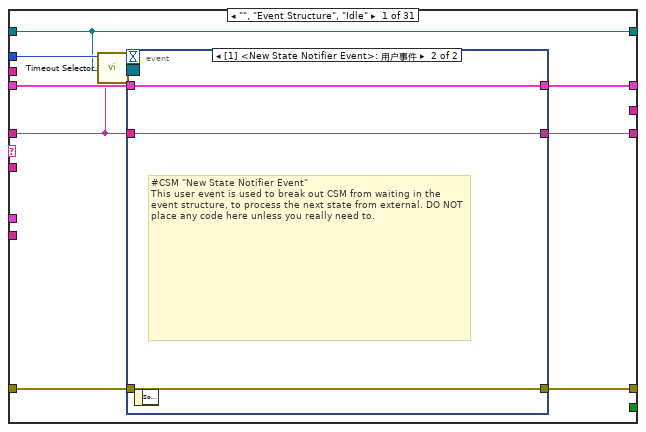
[diagram p2: hidden frame]
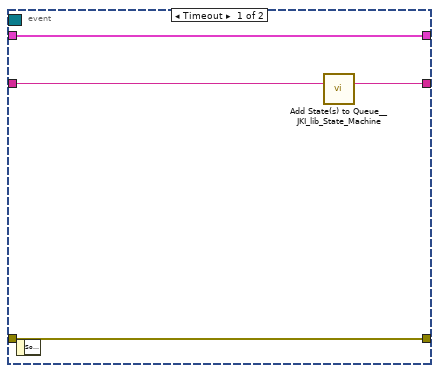
[diagram p3: hidden frame]
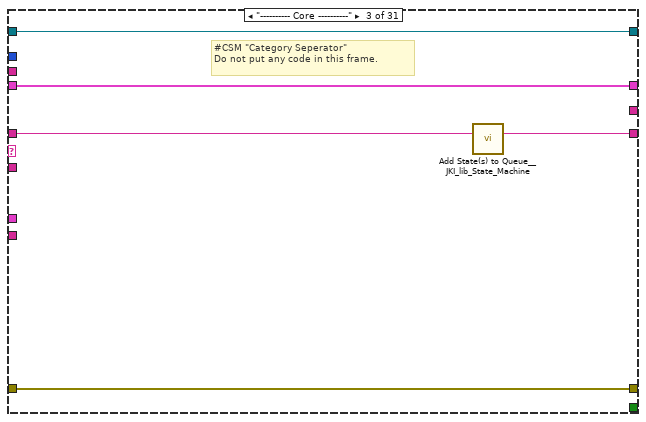
[diagram p5: hidden frame]
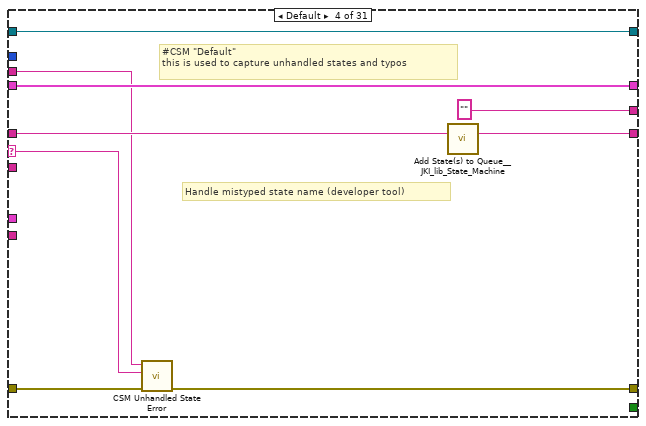
[diagram p6: hidden frame]
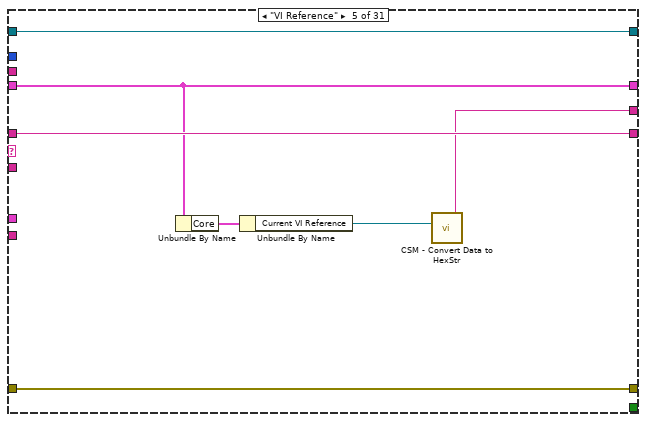
[diagram p7: hidden frame]
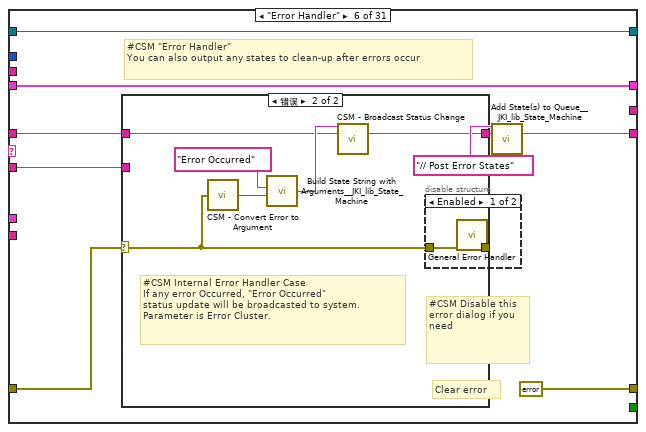
[diagram p8: hidden frame]
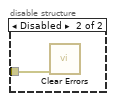
[diagram p9: hidden frame]
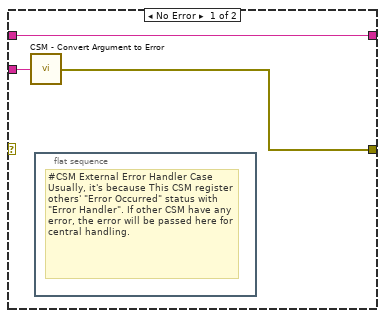
[diagram p10: hidden frame]
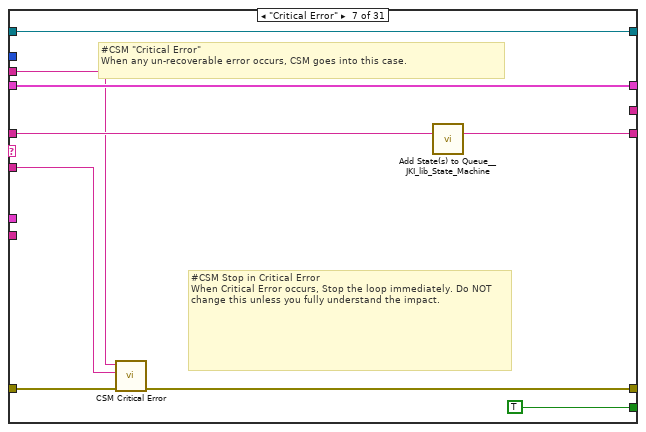
[diagram p11: hidden frame]
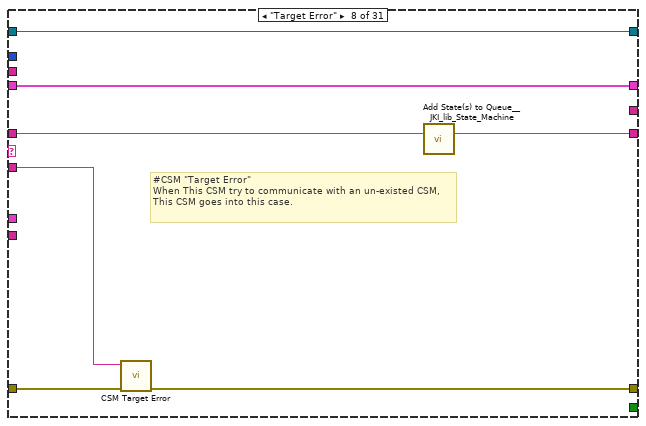
[diagram p12: hidden frame]
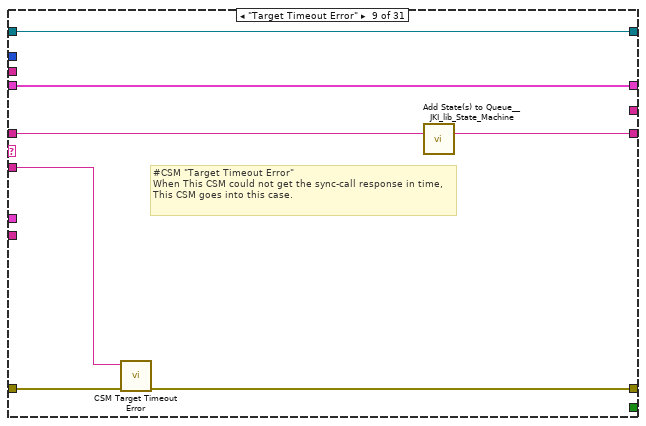
[diagram p13: hidden frame]
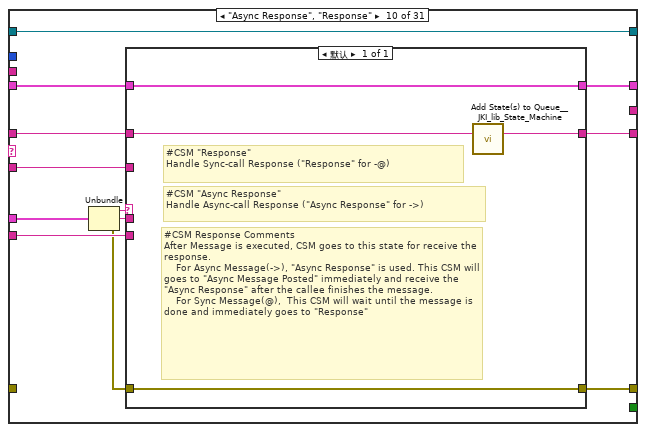
[diagram p14: hidden frame]
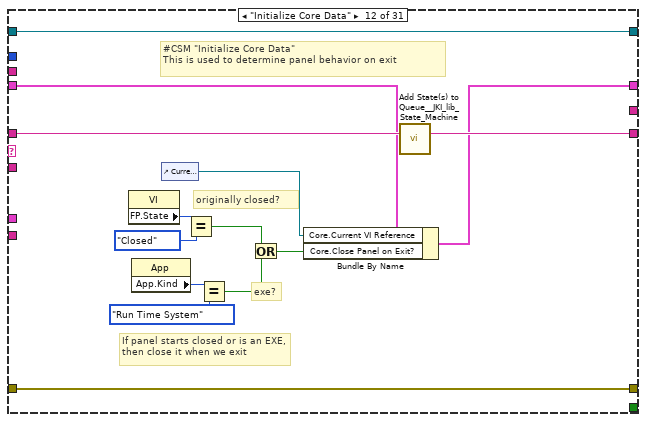
[diagram p16: hidden frame]
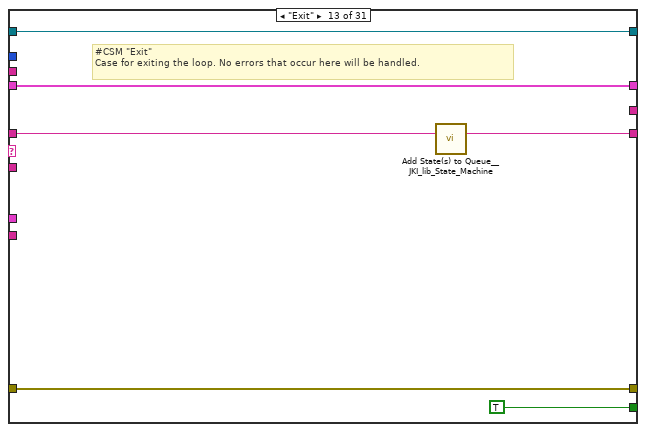
[diagram p17: hidden frame]
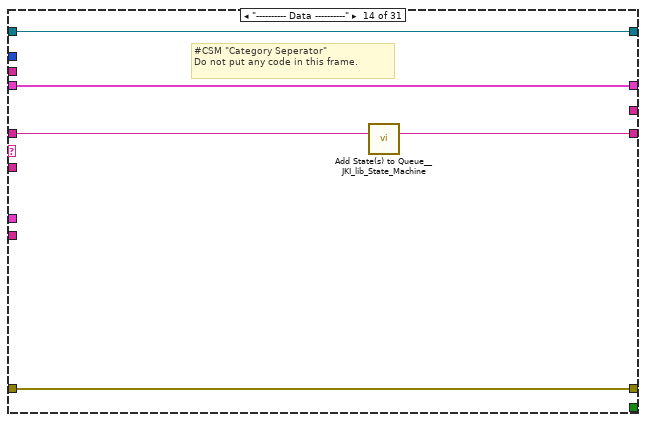
[diagram p18: hidden frame]
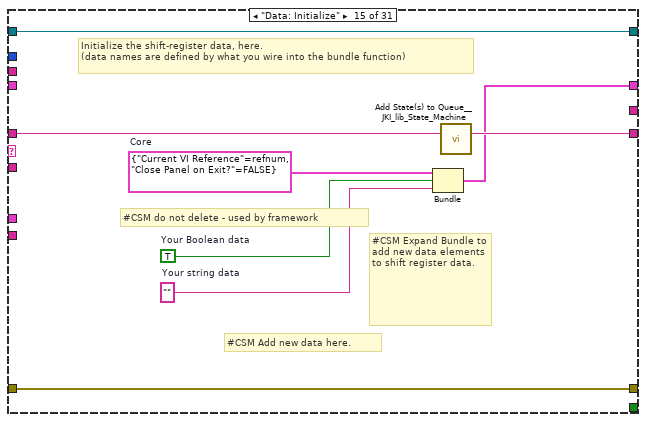
[diagram p19: hidden frame]
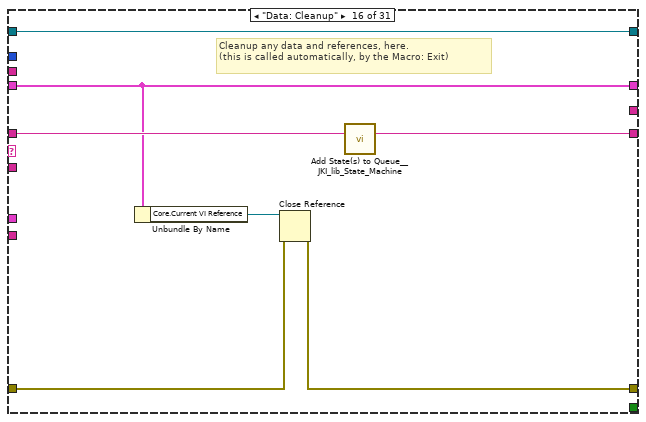
[diagram p20: hidden frame]
diagram:
  w14 = ""  # State
  # "to do：\n1. base cycle 小于0"
  # "Last Response Args"
  # "Internal Data"
  # "<< Internal Data"
  # "<< Response Args"
  # "<< Remaining States"
  # "Timeout to Send State(s) to CSM"
  # "Last Response Args"
  # "Internal Data"
  # "#CSM Name of the CSM\nIf you won't post any state from other CSM, leave this control blank."
  # "#CSM This controls the loop rate\nIt means wait forever until new message is coming"
  # "<< Internal Data"
  # "<< Response Args"
  # "<< Remaining States"
  n1 = case shown="False" "子程序？" {
    tunnel: [w16 errorcluster {"status"=FALSE, "code"=0, "source"=""} ("Error out")] -> w10
    frame False {
      n2 = call-poly <userlib>:"CSM - Read File Logger Configuration from INI String.vi"("Section Name(\"FileLogger\")"="FileLogger" ("Section Name(\"\" as Default)")) -> ("FileLogger Configuration-v1"=w23:T8)  [unwired: 7 in, 1 out]
      n3 = Unbundle By Name(w23) -> ("Enable"=w22:bool, "Limit"=w21:cluster{"FileSize":i64, "FileNum":i32}, "Timestamp.Format"=w19:string, "AutoExit"=w20:bool)
      n4 = call <vilib>:"Application Directory.vi"() -> ("Application Directory"=w28:path)
      n5 = Build Path(base path=w28, name or relative path="Blood Glucose System.csmlog") -> (appended path=w26:path)
      n6 = call <userlib>:"CSM - Start File Logger.vi"("Timestamp Format"=w19, "Log Limit"=w21, "Watchdog? (T)"=w22, "Exit When All Module Exist? (F)"=w20, "Log File Path"=w26) -> ("error out"=w25:errorcluster)  [unwired: 4 in, 2 out]
      n7 = call <userlib>:"CSM - Start Watchdog to Ensure All Modules Exit.vi"("error in (no error)"=w25) -> ("error out"=w17:errorcluster)  [unwired: 10 in]
      n8 = call <userlib>:"CSM - Config MassData Parameter Cache Size.vi"("Error in"=w17, "Size (50M)"=10000000 ("size(1M)")) -> ("Error out"=w16:errorcluster)  [unwired: 9 in]
    }
    frame True {
    }
  }
  n9 = call <vilib>:"Add State(s) to Queue__JKI_lib_State_Machine.vi"("State(s) in (\"\")"="Macro: Initialize" ("Init State(\"Macro: Initialize\")")) -> ("States Out"=w11:string)  [unwired: 14 in]
  n10 = while "Communicable State Machine(CSM) 2025" {
    shift-right: [w31] -> _
    shift-left: _ -> [w30]
    shift-right: [w45] -> w8
    shift-left: w10 -> [w34]
    shift-right: [w32] -> _
    shift-left: w11 -> [w46]
    tunnel: "CSM Name" -> [w41]
    shift-right: [w42] -> _
    shift-left: _ -> [w36]
    stop <- w44 stop-if-true
    w43 = -1  # TMO
    # "#CSM Debug State History\n(delete if unneeded)"
    # "-><interrupt>"
    # "-><status>"
    # "-><unregister>"
    # "-><register>"
    # "-@"
    # "->"
    # "->|"
    # "publish interrupt"
    # "publish status"
    # "Unregister Status"
    # "Register Status"
    # "Sync"
    # "Async with Reply"
    # "Async & No-Reply"
    # "JKI-SM Copyright © 2018 JKI - http://jki.net/state-machine CSM Copyright ?2025 NEVSTOP https://github.com/NEVSTOP-LAB"
    # "copy this to create labels for wires"
    # "System_Label"
    n11 = call <userlib>:"Parse State Queue++.vi"("State Queue"=w46, "Name (\"\" to Use UUID)"=w41, "Response Arguments"=w36, "Previous Error"=w34, "Dequeue (1 ms)"=w43) -> ("Name Used"=w35:string, "Remaining States"=w47:string, "Current State"=w37:string, "Arguments"=w38:string, "Additional Information"=w39:T15, "Source CSM"=w40:string)  [unwired: 5 in]
    n12 = call <userlib>:"CSM - Internal State Debug Log History.vi"("State"=w37, "Arguments (\"\")"=w38, ">> Response Source Message >>"=w39, "Source (\"\")"=w40) -> ("Debug Log"=→"State History":string)  [unwired: 11 in]
    n13 = case shown="\"UI: Initialize\"" w37 {
      selector: w37 -> [_ _ _ w58 _ _ _ _ _ _ _ _ _ _ _ _ _ _ _ _ _ _ _ _ _ _ _ _ _ _ _ _ _ _ _ _ _ _ _ _ _ _ _ _ _ _ _ w4195 w4226 w4257 _ _ w4342 w4355 w4368 w4382 w4391 _ w4426]
      tunnel: w47 -> [w48 w51 w54 w62 w67 w73 w98 w104 w110 w120 w127 w139 w143 w146 w162 w226 w242 w421 w424 w480 w493 w570 w600 w778 w1105 w1463 w1720 w2367 w2990 w3365 w3862 w3868 w3905 w3953 w3961 w3965 w3967 w3974 w3977 w4050 w4100 w4130 w4146 w4161 w4175 w4184 w4188 w4198 w4229 w4259 w4291 w4314 w4348 w4361 w4374 w4387 w4400 w4413 w4431]
      tunnel: w38 -> [_ _ _ _ _ w72 w94 w101 w107 w114 _ _ _ _ _ w224 _ _ _ _ _ _ _ _ _ _ _ _ _ _ _ _ w3897 _ _ _ _ _ w3979 w4016 _ _ _ w4155 _ w4183 _ _ _ _ _ _ w4344 w4357 w4370 w4384 w4396 _ w4428]
      tunnel: w30 -> [w49 w50 w52 w60 w66 w78 w96 w102 w108 w118 w126 w133 w141 w144 _ w170 w253 w416 w422 w427 w485 w560 w597 w735 w1061 w1425 w1643 w2365 w2940 w3378 w3860 w3866 w3883 w3951 w3959 w3964 w3969 w3976 w3995 w4052 w4074 w4132 w4140 w4152 w4166 w4181 w4190 w4192 w4224 w4254 w4287 w4304 w4339 w4353 w4366 w4380 w4394 w4405 w4418]
      tunnel: [_ _ _ w55 w68 errorcluster {"status"=FALSE, "code"=0, "source"=""} ("error out") w91 w99 w105 w121 _ _ _ _ _ _ w411 w417 _ _ w504 _ _ _ _ w1465 w1722 w2369 w2992 w3457 _ _ _ _ _ w3966 _ _ w3996 w4053 w4102 w4133 w4148 w4163 w4177 w4186 _ _ _ _ _ _ _ _ _ _ w4402 w4415 _] -> w45
      tunnel: w34 -> [_ _ _ w56 w68 w76 w92 w100 w106 _ _ _ _ _ _ _ w411 w418 _ _ w504 _ _ _ _ w1465 w1722 w2369 w2992 w3457 _ _ _ _ _ w3966 _ _ w3996 w4053 w4102 w4133 w4148 w4163 w4177 w4186 _ _ _ _ _ _ _ _ _ _ w4402 w4415 _]
      tunnel: [w48 w51 w53 w61 w67 w74 w97 w103 w109 w119 w127 w138 w142 w145 w161 w225 w243 w420 w423 w479 w494 w569 w599 w777 w1104 w1464 w1721 w2368 w2991 w3366 w3861 w3867 w3904 w3952 w3960 w3965 w3968 w3975 w3978 w4051 w4101 w4131 w4147 w4162 w4176 w4185 w4189 w4199 w4230 w4260 w4292 w4315 w4349 w4362 w4375 w4388 w4401 w4414 w4432] -> w32
      tunnel: [_ _ _ _ _ _ TRUE _ _ _ _ _ TRUE _ _ _ _ _ _ _ _ _ _ _ _ _ _ _ _ _ _ _ _ _ _ _ _ _ _ _ _ _ _ _ _ _ _ _ _ _ _ _ _ _ _ _ _ _ _] -> w44
      tunnel: [w49 w50 w52 w60 w66 w78 w96 w102 w108 w117 w126 w137 w141 w144 w160 w175 w253 w416 w422 w426 w486 w560 w597 w735 w1061 w1425 w1643 w2365 w2940 w3378 w3860 w3866 w3873 w3951 w3959 w3964 w3969 w3976 w3995 w4052 w4074 w4132 w4139 w4151 w4165 w4179 w4190 w4196 w4227 w4255 w4290 w4302 w4338 w4351 w4364 w4378 w4393 w4404 w4417] -> w31
      tunnel: w40 -> [_ _ _ _ _ w71 _ _ _ w115 _ _ _ _ _ _ _ _ _ _ _ _ _ _ _ _ _ _ _ _ _ _ _ _ _ _ _ _ _ _ _ _ _ _ _ _ _ _ _ _ _ _ _ _ _ _ _ _ _]
      tunnel: w39 -> [_ _ _ _ _ w70 _ _ _ w116 _ _ _ _ _ _ _ _ _ _ _ _ _ _ _ _ _ _ _ _ _ _ _ _ _ _ _ _ _ _ _ _ _ _ _ _ _ _ _ _ _ _ _ _ _ _ _ _ _]
      tunnel: [_ _ _ "" w63 _ _ _ _ _ _ _ _ _ _ _ _ _ _ _ _ _ _ _ _ _ _ _ _ _ _ _ _ _ _ _ _ _ _ _ _ _ _ _ _ _ _ _ _ _ _ _ _ _ _ _ _ _ _] -> w42
      tunnel: w35 -> [_ _ _ w57 _ _ w93 _ _ _ _ _ _ _ w147 w186 _ w414 _ w458 w490 _ _ _ _ _ _ _ _ _ _ w3864 _ w3949 w3957 _ _ _ _ _ _ _ _ _ _ _ _ w4197 w4228 w4258 _ _ w4346 w4359 w4372 w4386 w4398 w4409 w4430]
      frame "", "Idle" {
        # "#CSM \"Idle/Event Handler\"\nexecutes when the state queue is empty"
      }
      frame "CSM Documentation" {
        # "#CSM State Syntax\n\n// Comment line, all text to the right of “//” will be ignored\n// Local Message Example\nDoSth: DoA >> Arguments\n\n// Sync Call Example\nAPI: xxxx >> Arguments -@ TargetModule\n\n// Async Call Example\nAPI: xxxx >> Arguments -> TargetModule\n\n// Async Call without Reply Example\nAPI: xxxx >> Arguments ->| TargetModule\n\n// Broadcast normal status:\nStatus >> StatusArguments  -><status>\n\n// Broadcast Interrupt status:\nInterrupt >> StatusArguments  -><interrupt>\n\n// Register Source Module's status to Handler Module\nStatus@Source Module >> Handler Module@Handler Module -><register>\n\n// Unegister Source Module's status\nStatus@Source Module >> Handler Module -><unregister>"
        # "#CSM README FIRST\n\nCommunicable State Machine(CSM) is a LabVIEW application framework that builds upon JKI State Machine(JKISM). It follows the pattern of JKISM and extends the keywords to describe message communication between modules, including concepts such as Sync-Message, Async-Message, Subscription/Unsubscription of status - essential elements for creating reusable code modules. For more information, please visit the CSM wiki: https://nevstop-lab.github.io/CSM-Wiki/\n\nFor instructions on JKI State Machine, visit: \n    http://jki.net/state-machine/\nFor information about CSM, visit: \n    https://github.com/NEVSTOP-LAB"
        # "#CSM \"Documentation\"\nCase for holding CSM Documenation"
      }
      frame "---------- Core ----------" {
        # "#CSM \"Category Seperator\"\nDo not put any code in this frame."
        n14 = call <vilib>:"Add State(s) to Queue__JKI_lib_State_Machine.vi"("State(s) in (\"\")"=w54) -> ("States Out"=w53:string)  [unwired: 14 in]
      }
      frame Default {
        # "#CSM \"Default\"\nthis is used to capture unhandled states and typos"
        n15 = call <userlib>:"CSM Unhandled State Error.vi"("error in (no error)"=w56, "Undefined State"=w58, "CSM Name"=w57) -> ("error out"=w55:errorcluster)  [unwired: 8 in]
        n16 = call <vilib>:"Add State(s) to Queue__JKI_lib_State_Machine.vi"("State(s) in (\"\")"=w62) -> ("States Out"=w61:string)  [unwired: 14 in]
      }
      frame "VI Reference" {
        n17 = Unbundle By Name(w66) -> ("Core"=w65:T16)
        n18 = Unbundle By Name(w65) -> ("Current VI Reference"=w64:refnum<vi>)
        n19 = call <userlib>:"CSM - Convert Data to HexStr.vi"("Variant"=w64) -> ("HEX String (0-9,A-F)"=w63:string)  [unwired: 8 in]
      }
      frame "Error Handler" {
        # "#CSM \"Error Handler\"\nYou can also output any states to clean-up after errors occur"
        # "Clear error"
        n20 = case shown="错误" w76 {
          selector: w76 -> [_ w85]
          tunnel: [w83 w87] -> w75
          tunnel: w73 -> [w83 w86]
          tunnel: w72 -> [w82 _]
          tunnel: w71 -> [_ _]
          tunnel: w70 -> [_ _]
          tunnel: [w80 w85] -> w69
          frame No Error {
            n21 = call <userlib>:"CSM - Convert Argument to Error.vi"("Argument"=w82) -> ("Error"=w81:errorcluster)  [unwired: 4 in]
            n22 = flat-sequence {
              tunnel: w81 -> [w84]
              tunnel: [w84] -> w80
              frame #0 {
              }
            }
          }
          frame Error {
            # "#CSM Internal Error Handler Case \nIf any error Occurred, \"Error Occurred\" \nstatus update will be broadcasted to system.\nParameter is Error Cluster."
            n23 = call <userlib>:"CSM - Convert Error to Argument.vi"("Error"=w85) -> ("Argument"=w89:string)  [unwired: 4 in]
            n24 = call <vilib>:"Build State String with Arguments__JKI_lib_State_Machine.vi"("Arguments (\"\")"=w89, "State"="Error Occurred" ("Status with Arguments")) -> ("State with Arguments"=w88:string)  [unwired: 4 in]
            n25 = call <userlib>:"CSM - Broadcast Status Change.vi"("Status With Arguments"=w88, "State Queue"=w86) -> ("Remaining States"=w87:string)  [unwired: 13 in]
          }
        }
        "Error Occurred" <- w69
        n26 = call <vilib>:"Add State(s) to Queue__JKI_lib_State_Machine.vi"("State(s) in Front (\"\")"="// Post Error States", "State(s) in (\"\")"=w75) -> ("States Out"=w74:string)  [unwired: 13 in]
      }
      frame "Critical Error" {
        # "#CSM \"Critical Error\"\nWhen any un-recoverable error occurs, CSM goes into this case."
        # "#CSM Stop in Critical Error\nWhen Critical Error occurs, Stop the loop immediately. Do NOT change this unless you fully understand the impact."
        n27 = call <userlib>:"CSM Critical Error.vi"("error in (no error)"=w92, "Arugments (As Reason)"=w94, "CSM Name"=w93) -> ("error out"=w91:errorcluster)  [unwired: 8 in]
        n28 = call <vilib>:"Add State(s) to Queue__JKI_lib_State_Machine.vi"("State(s) in (\"\")"=w98) -> ("States Out"=w97:string)  [unwired: 14 in]
      }
      frame "Target Timeout Error" {
        # "#CSM \"Target Timeout Error\"\nWhen This CSM could not get the sync-call response in time, This CSM goes into this case."
        n29 = call <userlib>:"CSM Target Timeout Error.vi"("error in (no error)"=w100, "Arguments (As CSM Name)"=w101) -> ("error out"=w99:errorcluster)  [unwired: 9 in]
        n30 = call <vilib>:"Add State(s) to Queue__JKI_lib_State_Machine.vi"("State(s) in (\"\")"=w104) -> ("States Out"=w103:string)  [unwired: 14 in]
      }
      frame "Target Error" {
        # "#CSM \"Target Error\"\nWhen This CSM try to communicate with an un-existed CSM, This CSM goes into this case."
        n31 = call <userlib>:"CSM Target Error.vi"("error in (no error)"=w106, "Arguments (As CSM Name)"=w107) -> ("error out"=w105:errorcluster)  [unwired: 9 in]
        n32 = call <vilib>:"Add State(s) to Queue__JKI_lib_State_Machine.vi"("State(s) in (\"\")"=w110) -> ("States Out"=w109:string)  [unwired: 14 in]
      }
      frame "Async Response", "Response" {
        n33 = Unbundle(w116) -> ("‘State"=w113:string, "’Arguments"=w112:string, "’Error"=w111:errorcluster)
        n34 = case shown="默认" w113 {
          tunnel: [w122] -> w119
          tunnel: w120 -> [w123]
          tunnel: [w125] -> w117
          tunnel: w118 -> [w125]
          tunnel: [w124] -> w121
          tunnel: w111 -> [w124]
          tunnel: w115 -> [_]
          tunnel: w114 -> [_]
          tunnel: w112 -> [_]
          frame 默认 {
            # "#CSM \"Async Response\"\nHandle Async-call Response (\"Async Response\" for ->)"
            # "#CSM \"Response\"\nHandle Sync-call Response (\"Response\" for -@)"
            # "#CSM Response Comments\nAfter Message is executed, CSM goes to this state for receive the response.\n    For Async Message(->), \"Async Response\" is used. This CSM will goes to \"Async Message Posted\" immediately and receive the \"Async Response\" after the callee finishes the message.\n    For Sync Message(@),  This CSM will wait until the message is done and immediately goes to \"Response\""
            n35 = call <vilib>:"Add State(s) to Queue__JKI_lib_State_Machine.vi"("State(s) in (\"\")"=w123) -> ("States Out"=w122:string)  [unwired: 14 in]
          }
        }
      }
      frame "Async Message Posted" {
        # "#CSM \"Async Message Posted\"\nAfter Async Message is posted (-> or ->| ), CSM goes to this state for post-action.\nYou can use Argument - State to tell which Async Message is called."
      }
      frame "Initialize Core Data" {
        # "#CSM \"Initialize Core Data\"\nThis is used to determine panel behavior on exit"
        # "originally closed?"
        # "exe?"
        # "If panel starts closed or is an EXE, then close it when we exit"
        n36 = property class="VI"() -> ("FP.State"=w130:T9)  [unwired: 2 in, 2 out]
        n37 = property class="App"() -> ("App.Kind"=w136:T10)  [unwired: 2 in, 2 out]
        n38 = control-ref of="Current VI Reference"() -> (w131:refnum<vi>)
        n39 = Equal?(x=w130, y=T9."Closed" ("Front Panel Window:State")) -> (x = y?=w128:bool)
        n40 = Equal?(x=w136, y=T10."Run Time System" ("Application:Kind")) -> (x = y?=w134:bool)
        n41 = Or(x=w128, y=w134) -> (x .or. y?=w132:bool)
        n42 = call <vilib>:"Add State(s) to Queue__JKI_lib_State_Machine.vi"("State(s) in (\"\")"=w139) -> ("States Out"=w138:string)  [unwired: 14 in]
        n43 = Bundle By Name(cluster=w133, "Core.Current VI Reference"=w131, "Core.Close Panel on Exit?"=w132) -> (w137:T20)
      }
      frame "Exit" {
        # "#CSM \"Exit\"\nCase for exiting the loop. No errors that occur here will be handled."
        n44 = call <vilib>:"Add State(s) to Queue__JKI_lib_State_Machine.vi"("State(s) in (\"\")"=w143) -> ("States Out"=w142:string)  [unwired: 14 in]
      }
      frame "---------- Data ----------" {
        # "#CSM \"Category Seperator\"\nDo not put any code in this frame."
        n45 = call <vilib>:"Add State(s) to Queue__JKI_lib_State_Machine.vi"("State(s) in (\"\")"=w146) -> ("States Out"=w145:string)  [unwired: 14 in]
      }
      frame "Data: Initialize" {
        w149 = T19 {"控制"={"信号采集设备和供电"="Dev1", "自动停止(周期)"=inf, "自动停止(时间, min)"=inf, "测头类型"=enum."5环-单测头", "测量波长"=[]}, "校准"={"温度校准值（每度）"=[[0.0, 0.0, 0.0, 0.0, 0.0, 0.0, 0.00013, 0.00013, 0.00013, 0.00013, 0.00013, 0.00013], [0.0, 0.0, 0.0, 0.0, 0.0, 0.0, 0.00013, 0.00013, 0.00013, 0.00013, 0.00013, 0.00013], [0.0, 0.0, 0.0, 0.0, 0.0, 0.0, 0.00013, 0.00013, 0.00013, 0.00013, 0.00013, 0.00013], [0.0, 0.0, 0.0, 0.0, 0.0, 0.0, 0.00013, 0.00013, 0.00013, 0.00013, 0.00013, 0.00013], [0.0, 0.0, 0.0, 0.0, 0.0, 0.0, 0.00013, 0.00013, 0.00013, 0.00013, 0.00013, 0.00013], [0.0, 0.0, 0.0, 0.0, 0.0, 0.0, 0.00013, 0.00013, 0.00013, 0.00013, 0.00013, 0.00013], [0.0, 0.0, 0.0, 0.0, 0.0, 0.0, 0.00013, 0.00013, 0.00013, 0.00013, 0.00013, 0.00013], [0.0, 0.0, 0.0, 0.0, 0.0, 0.0, 0.00013, 0.00013, 0.00013, 0.00013, 0.00013, 0.00013], [0.0, 0.0, 0.0, 0.0, 0.0, 0.0, 0.00013, 0.00013, 0.00013, 0.00013, 0.00013, 0.00013], [0.0, 0.0, 0.0, 0.0, 0.0, 0.0, 0.00013, 0.00013, 0.00013, 0.00013, 0.00013, 0.00013], [0.00013, 0.00013, 0.00013, 0.00013, 0.00013, 0.00013, 0.00013, 0.00013, 0.00013, 0.00013, 0.00013, 0.00013], [0.00013, 0.00013, 0.00013, 0.00013, 0.00013, 0.00013, 0.00013, 0.00013, 0.00013, 0.00013, 0.00013, 0.00013], [0.00013, 0.00013, 0.00013, 0.00013, 0.00013, 0.00013, 0.00013, 0.00013, 0.00013, 0.00013, 0.00013, 0.00013], [0.00013, 0.00013, 0.00013, 0.00013, 0.00013, 0.00013, 0.00013, 0.00013, 0.00013, 0.00013, 0.00013, 0.00013], [0.00013, 0.00013, 0.00013, 0.00013, 0.00013, 0.00013, 0.00013, 0.00013, 0.00013, 0.00013, 0.00013, 0.00013], [0.00013, 0.00013, 0.00013, 0.00013, 0.00013, 0.00013, 0.00013, 0.00013, 0.00013, 0.00013, 0.00013, 0.00013], [0.00013, 0.00013, 0.00013, 0.00013, 0.00013, 0.00013, 0.00013, 0.00013, 0.00013, 0.00013, 0.00013, 0.00013], [0.00013, 0.00013, 0.00013, 0.00013, 0.00013, 0.00013, 0.00013, 0.00013, 0.00013, 0.00013, 0.00013, 0.00013], [0.00013, 0.00013, 0.00013, 0.00013, 0.00013, 0.00013, 0.00013, 0.00013, 0.00013, 0.00013, 0.00013, 0.00013], [0.00013, 0.00013, 0.00013, 0.00013, 0.00013, 0.00013, 0.00013, 0.00013, 0.00013, 0.00013, 0.00013, 0.00013]], "温度校准通道"=enum."温度通道2"}, "图表相关"={"分段颜色"=enum."蓝色", "程序开始时间"=timestamp(0 s since 1904-01-01), "基准索引"=0}, "Save Delay"={"放下周期"=0, "进度"=enum."拿起"}, "波长差分"={"X"=4, "Y"=0, "差分X"=9, "差分Y"=9, "k"=1.0, "X2"=4, "Y2"=0, "差分X2"=7, "差分Y2"=7, "k2"=1.0, "X3"=4, "Y3"=0, "差分X3"=8, "差分Y3"=8, "k3"=1.0}}  # Indicators
        w157 = T18 {"采集时间"=timestamp(0 s since 1904-01-01), "采集时间(dbl)"=0.0, "Data"=[0.0, 0.0, 0.0, 0.0, 0.0, 0.0, 0.0], "当前运行信息"={"当前周期"=0, "当前次数"=0, "测量周期"=0, "当前索引子集"=[], "当前波长"=0}, "暗电流校准值"=[], "Logging Settings"={"是否保存？"=FALSE, "波长结束？"=FALSE, "周期结束？"=FALSE}, "原始值"={"1环(原始值)"=[], "2环(原始值)"=[], "3环(原始值)"=[], "4环(原始值)"=[], "5环(原始值)"=[], "6环(原始值)"=[], "7环(原始值)"=[]}, "校准值"={"1环(校准值)"=[], "2环(校准值)"=[], "3环(校准值)"=[], "4环(校准值)"=[], "5环(校准值)"=[], "6环(校准值)"=[], "7环(校准值)"=[]}}  # Time and Data
        w154 = T17 {"设备信息"={"初始索引子集"=[], "模拟信号采集通道"="Dev1", "数字-供电"="", "数字-光控"="", "光控设备"="", "光电设备分离？"=FALSE, "光谱保存路径"=path "", "环数"=0}, "测量控制"={"测头拿起"=FALSE, "起始保存"=FALSE, "测头供电"=TRUE, "测头出光"=TRUE}, "测量"={"每波长测量次数"=5, "波长"=[0, 0, 0, 0, 0, 0], "起始周期"=0, "起始测量周期"=0}, "等待"={"等待时间(s)"=0.0, "等待方式"=FALSE, "每x周期/点等待"=8, "等待时"=enum."无电无光"}, "校准"={"暗电流校准值初值"=[], "温度校准值"=[0.0, 0.0, 0.0, 0.0, 0.0, 0.0, 0.00013, 0.00013, 0.00013, 0.00013, 0.00013, 0.00013], "校准模式"=enum."逐周期"}, "图表相关"={"文件-时间"=""}, "CSM"={"CSM Name"=""}}  # Sample Settings
        w159 = T16 {"Current VI Reference"=refnum, "Close Panel on Exit?"=FALSE}  # Core
        # "#CSM \"Data: Initialize\"\nInitialize the shift-register data, here.\n(data names are defined by what you wire into the bundle function)"
        # "#CSM do not delete - used by framework"
        # "#CSM Data names and types of shift register data are defined by this bundle."
        n46 = local read "子程序？"() -> (w156:bool)
        n47 = call "CSM - Read Cluster Elements From Session.vim"("Section Name (\"\" as Default)"=w147, "Cluster"=w154) -> ("Cluster out"=w155:T17)  [unwired: 6 in, 1 out]
        n48 = call "CSM - Read Cluster Elements From Session.vim"("Section Name (\"\" as Default)"=w147, "Cluster"=w149) -> ("Cluster out"=w150:T19)  [unwired: 6 in, 1 out]
        n49 = Select(t=w155, s=TRUE, f=w154) -> (s? t:f=w152:T17)
        n50 = Select(t=w150, s=TRUE, f=w149) -> (s? t:f=w148:T19)
        n51 = local write "Error Occurred"(errorcluster {"status"=FALSE, "code"=0, "source"=""} ("Error Occurred")) -> ()
        n52 = Bundle("Core"=w159, "Sample Settings"=w152, "Time and Data"=w157, "Indicators"=w148, "子程序？"=w156) -> (w160:T20)  [unwired: 1 in]
        n53 = call <vilib>:"Add State(s) to Queue__JKI_lib_State_Machine.vi"("State(s) in (\"\")"=w162) -> ("States Out"=w161:string)  [unwired: 14 in]
      }
      frame "Data: Update Indicators" {
        w223 = T18 {"采集时间"=timestamp(0 s since 1904-01-01), "采集时间(dbl)"=0.0, "Data"=[], "当前运行信息"={"当前周期"=0, "当前次数"=0, "测量周期"=0, "当前索引子集"=[], "当前波长"=0}, "暗电流校准值"=[], "Logging Settings"={"是否保存？"=FALSE, "波长结束？"=FALSE, "周期结束？"=FALSE}, "原始值"={"1环(原始值)"=[], "2环(原始值)"=[], "3环(原始值)"=[], "4环(原始值)"=[], "5环(原始值)"=[], "6环(原始值)"=[], "7环(原始值)"=[]}, "校准值"={"1环(校准值)"=[], "2环(校准值)"=[], "3环(校准值)"=[], "4环(校准值)"=[], "5环(校准值)"=[], "6环(校准值)"=[], "7环(校准值)"=[]}}  # Time and Data
        n54 = global read "辅助系统全局变量 - T1.vi" "温度相关数据"() -> (w197:T21)
        n55 = Unbundle By Name(w197) -> ("温度采集"=w199:dbl[], "温度控制"=w200:dbl[], "压力测量"=w201:dbl[], "Zolix"=w202:dbl[], "步进电机"=w203:dbl[], "湿度测量"=w204:dbl[])
        n56 = local read "分段颜色"() -> (w184:enum32{"蓝色", "红色"})
        n57 = Decrement(x="校准通道") -> (x-1=w196:T6)
        n58 = local write "程序状态"("测量中" ("程序状态")) -> ()
        n59 = Build Array (concatenate)(w199, w200, w201, w202, w203, w204) -> (w198:dbl[])
        n60 = Index Array(array=w198, index=w196) -> (element=w195:dbl)
        "校准温度" <- w195
        n61 = call "CSM - Convert Argument to MassData.vim"("Type"=w223, "MassData Argument"=w224) -> ("Data"=w171:T18)  [unwired: 6 in, 1 out]
        n62 = Unbundle By Name(w170) -> ("Sample Settings.测量.波长"=w189:i32[], "Sample Settings.测量.每波长测量次数"=w165:i32, "Indicators.校准.温度校准值（每度）"=w207:dbl[][], "Sample Settings.设备信息.光谱保存路径"=w191:path, "Sample Settings.图表相关.文件-时间"=w190:string, "Sample Settings.设备信息.初始索引子集"=w182:i8[])
        n63 = call "CSM Get Module Attribute.vim"("CSM Name"=w186, "Attribute"="分段颜色", "Default Value (Empty Variant)"=w184) -> ("Value"=w174:enum32{"蓝色", "红色"})  [unwired: 8 in, 4 out]
        n64 = Unbundle By Name(w171) -> ("暗电流校准值"=w172:dbl[], "Data"=w222:dbl[], "当前运行信息.当前周期"=w187:i32, "当前运行信息.当前次数"=→"第N次测量":i32, "当前运行信息.测量周期"=w166:i32, "当前运行信息.当前索引子集"=w194:i8[], "Logging Settings.波长结束？"=w178:bool, "Logging Settings.是否保存？"=w183:bool)
        "当前周期" <- w187
        "测量周期" <- w166
        n65 = call "CSM Set Module Attribute.vim"("CSM Name"=w186, "Attribute"="当前周期", "Value"=w187) -> ()  [unwired: 9 in, 4 out]
        n66 = local write "分段颜色"(w174) -> ()
        n67 = local write "是否保存"(w183) -> ()
        n68 = Index Array(array=w194) -> (element=w181:i8)  [unwired: 1 in]
        n69 = Index Array(array=w182, index=1 ("索引")) -> (element=w180:i8)
        n70 = Index Array(array=w189, index=w181) -> (element=→"当前波长":i32)
        n71 = Equal?(x=w181, y=w180) -> (x = y?=w179:bool)
        n72 = Multiply(x=w166, y=w165) -> (x*y=→"测量点数(图表)":i32)
        n73 = Index Array(array=w222) -> (element #1=→"1环":dbl, element #2=→"2环":dbl, element #3=→"3环":dbl, element #4=→"4环":dbl, element #5=→"5环":dbl, element #6=→"6环":dbl, element #7=→"7环":dbl)  [unwired: 7 in]
        n74 = Select(t=w207, s="是否校准？", f=dbl[][] []) -> (s? t:f=w211:dbl[][])
        n75 = local write "暗电流校准值"(w172) -> ()
        n76 = Subtract(x=w195, y="基准温度") -> (x-y=w212:dbl)
        n77 = Multiply(x=w212, y=w211) -> (x*y=w206:dbl[][])
        n78 = Index Array(array=w206, index (col)=w181) -> (element=w173:dbl[])  [unwired: 1 in]
        n79 = Compound Arithmetic op=AND(w179, w178) -> (w177:bool)
        n80 = Decrement(x=w166) -> (x-1=w168:i32)
        n81 = case shown="True" w177 {
          tunnel: w191 -> [_ w235]
          tunnel: w190 -> [_ w234]
          frame False {
          }
          frame True {
            n82 = Concatenate Strings(w234, "(校准后)-1环.dat" ("字符串")) -> (w238:string)
            n83 = Build Path(base path=w235, name or relative path=w238) -> (appended path=w236:path)
            n84 = call "数据保存判断.vi"("appended path"=w236) -> ("数据保存中?"=→"数据保存中？":bool)  [unwired: 10 in]
          }
        }
        n85 = Max & Min(x="A | Ad\n基准周期", y=w168) -> (min(x,y)=w169:i32)  [unwired: 1 out]
        n86 = Multiply(x=w169, y=w165) -> (x*y=w167:i32)
        n87 = Decrement(x=w167) -> (x-1=w164:i32)
        n88 = in-place {
          in-place-border: w174 -> [w232]
          in-place-border: w173 -> [w231]
          in-place-border: w172 -> [w230]
          in-place-border: w171 -> [w229]
          in-place-border: w164 -> [w228]
          n89 = in-place-cluster #1(w170) -> ()  [unwired: 5 out]
          n90 = in-place-cluster #1("Time and Data"=w229, "Sample Settings.校准.暗电流校准值初值"=w230, "Sample Settings.校准.温度校准值"=w231, "Indicators.图表相关.分段颜色"=w232, "Indicators.图表相关.基准索引"=w228) -> (w175:T20)
        }
        n91 = call <vilib>:"Add State(s) to Queue__JKI_lib_State_Machine.vi"("State(s) in Front (\"\")"="UI: Update Graph" ("State(s) in Front (\"\")"), "State(s) in (\"\")"=w226) -> ("States Out"=w225:string)  [unwired: 13 in]
      }
      frame "Data: Update SNR" {
        w327 = 1 ("索引")
        # "信噪比计算"
        n92 = Unbundle By Name(w253) -> ("Sample Settings.测量.波长"=w240:i32[], "Sample Settings.测量.每波长测量次数"=w252:i32, "Time and Data.当前运行信息.当前索引子集"=w251:i8[], "Time and Data.校准值.1环(校准值)"=w250:dbl[][], "Time and Data.校准值.2环(校准值)"=w249:dbl[][], "Time and Data.校准值.3环(校准值)"=w248:dbl[][], "Time and Data.校准值.4环(校准值)"=w247:dbl[][], "Time and Data.校准值.5环(校准值)"=w246:dbl[][], "Time and Data.校准值.6环(校准值)"=w245:dbl[][], "Time and Data.校准值.7环(校准值)"=w244:dbl[][])
        n93 = Reverse 1D Array(array=w251) -> (reversed array=w254:i8[])
        n94 = Subtract(x=w252, y=w327) -> (x-y=w328:i32)
        n95 = Index Array(array=w254) -> (element=w241:i8)  [unwired: 1 in]
        n96 = Array Subset(array=w250, index (col)=w327, length (col)=w328) -> (w402:dbl[][])  [unwired: 2 in]
        n97 = Array Subset(array=w249, index (col)=w327, length (col)=w328) -> (w401:dbl[][])  [unwired: 2 in]
        n98 = Array Subset(array=w248, index (col)=w327, length (col)=w328) -> (w400:dbl[][])  [unwired: 2 in]
        n99 = Array Subset(array=w247, index (col)=w327, length (col)=w328) -> (w399:dbl[][])  [unwired: 2 in]
        n100 = Array Subset(array=w246, index (col)=w327, length (col)=w328) -> (w372:dbl[][])  [unwired: 2 in]
        n101 = Array Subset(array=w245, index (col)=w327, length (col)=w328) -> (w330:dbl[][])  [unwired: 2 in]
        n102 = Array Subset(array=w244, index (col)=w327, length (col)=w328) -> (w329:dbl[][])  [unwired: 2 in]
        n103 = Index Array(array=w402, index (row)=w241) -> (element=w349:dbl[])  [unwired: 1 in]
        n104 = Index Array(array=w401, index (row)=w241) -> (element=w350:dbl[])  [unwired: 1 in]
        n105 = Index Array(array=w400, index (row)=w241) -> (element=w351:dbl[])  [unwired: 1 in]
        n106 = Index Array(array=w399, index (row)=w241) -> (element=w352:dbl[])  [unwired: 1 in]
        n107 = Index Array(array=w372, index (row)=w241) -> (element=w353:dbl[])  [unwired: 1 in]
        n108 = Index Array(array=w330, index (row)=w241) -> (element=w265:dbl[])  [unwired: 1 in]
        n109 = Index Array(array=w329, index (row)=w241) -> (element=w264:dbl[])  [unwired: 1 in]
        n110 = Natural Logarithm(1:w264) -> (0:w257:dbl[])
        n111 = Natural Logarithm(1:w265) -> (0:w258:dbl[])
        n112 = Index Array(array=w240, index=w241) -> (element=→"波长":i32)
        n113 = Natural Logarithm(1:w353) -> (0:w259:dbl[])
        n114 = Natural Logarithm(1:w352) -> (0:w260:dbl[])
        n115 = Natural Logarithm(1:w351) -> (0:w261:dbl[])
        n116 = Natural Logarithm(1:w350) -> (0:w262:dbl[])
        n117 = Natural Logarithm(1:w349) -> (0:w263:dbl[])
        n118 = Subtract(x=w263, y=w262) -> (x-y=w381:dbl[])
        n119 = Subtract(x=w263, y=w261) -> (x-y=w373:dbl[])
        n120 = Subtract(x=w263, y=w260) -> (x-y=w365:dbl[])
        n121 = Subtract(x=w263, y=w259) -> (x-y=w367:dbl[])
        n122 = Subtract(x=w262, y=w261) -> (x-y=w394:dbl[])
        n123 = Subtract(x=w262, y=w260) -> (x-y=w391:dbl[])
        n124 = Subtract(x=w262, y=w259) -> (x-y=w388:dbl[])
        n125 = Subtract(x=w261, y=w260) -> (x-y=w361:dbl[])
        n126 = Subtract(x=w261, y=w259) -> (x-y=w358:dbl[])
        n127 = Subtract(x=w260, y=w259) -> (x-y=w332:dbl[])
        n128 = Subtract(x=w263, y=w258) -> (x-y=w306:dbl[])
        n129 = Subtract(x=w263, y=w257) -> (x-y=w298:dbl[])
        n130 = Subtract(x=w262, y=w258) -> (x-y=w294:dbl[])
        n131 = Subtract(x=w262, y=w257) -> (x-y=w296:dbl[])
        n132 = Subtract(x=w261, y=w258) -> (x-y=w319:dbl[])
        n133 = Subtract(x=w261, y=w257) -> (x-y=w316:dbl[])
        n134 = Subtract(x=w260, y=w258) -> (x-y=w313:dbl[])
        n135 = Subtract(x=w260, y=w257) -> (x-y=w290:dbl[])
        n136 = Subtract(x=w259, y=w258) -> (x-y=w287:dbl[])
        n137 = Subtract(x=w259, y=w257) -> (x-y=w282:dbl[])
        n138 = Subtract(x=w258, y=w257) -> (x-y=w279:dbl[])
        n139 = call <vilib>:"Std Deviation and Variance.vi"("X"=w349) -> ("mean"=w409:dbl, "standard deviation"=w410:dbl)  [unwired: 1 in, 1 out]
        n140 = call <vilib>:"Std Deviation and Variance.vi"("X"=w350) -> ("mean"=w408:dbl, "standard deviation"=w407:dbl)  [unwired: 1 in, 1 out]
        n141 = call <vilib>:"Std Deviation and Variance.vi"("X"=w351) -> ("mean"=w405:dbl, "standard deviation"=w406:dbl)  [unwired: 1 in, 1 out]
        n142 = call <vilib>:"Std Deviation and Variance.vi"("X"=w352) -> ("mean"=w404:dbl, "standard deviation"=w403:dbl)  [unwired: 1 in, 1 out]
        n143 = call <vilib>:"Std Deviation and Variance.vi"("X"=w353) -> ("mean"=w369:dbl, "standard deviation"=w370:dbl)  [unwired: 1 in, 1 out]
        n144 = call <vilib>:"Std Deviation and Variance.vi"("X"=w265) -> ("mean"=w324:dbl, "standard deviation"=w325:dbl)  [unwired: 1 in, 1 out]
        n145 = call <vilib>:"Std Deviation and Variance.vi"("X"=w264) -> ("mean"=w321:dbl, "standard deviation"=w322:dbl)  [unwired: 1 in, 1 out]
        n146 = call <vilib>:"Std Deviation and Variance.vi"("X"=w381) -> ("mean"=w382:dbl, "standard deviation"=w380:dbl)  [unwired: 1 in, 1 out]
        n147 = call <vilib>:"Std Deviation and Variance.vi"("X"=w373) -> ("mean"=w378:dbl, "standard deviation"=w379:dbl)  [unwired: 1 in, 1 out]
        n148 = call <vilib>:"Std Deviation and Variance.vi"("X"=w365) -> ("mean"=w375:dbl, "standard deviation"=w374:dbl)  [unwired: 1 in, 1 out]
        n149 = call <vilib>:"Std Deviation and Variance.vi"("X"=w367) -> ("mean"=w366:dbl, "standard deviation"=w368:dbl)  [unwired: 1 in, 1 out]
        n150 = call <vilib>:"Std Deviation and Variance.vi"("X"=w394) -> ("mean"=w393:dbl, "standard deviation"=w395:dbl)  [unwired: 1 in, 1 out]
        n151 = call <vilib>:"Std Deviation and Variance.vi"("X"=w391) -> ("mean"=w392:dbl, "standard deviation"=w390:dbl)  [unwired: 1 in, 1 out]
        n152 = call <vilib>:"Std Deviation and Variance.vi"("X"=w388) -> ("mean"=w387:dbl, "standard deviation"=w389:dbl)  [unwired: 1 in, 1 out]
        n153 = call <vilib>:"Std Deviation and Variance.vi"("X"=w361) -> ("mean"=w362:dbl, "standard deviation"=w360:dbl)  [unwired: 1 in, 1 out]
        n154 = call <vilib>:"Std Deviation and Variance.vi"("X"=w358) -> ("mean"=w357:dbl, "standard deviation"=w359:dbl)  [unwired: 1 in, 1 out]
        n155 = call <vilib>:"Std Deviation and Variance.vi"("X"=w332) -> ("mean"=w331:dbl, "standard deviation"=w354:dbl)  [unwired: 1 in, 1 out]
        n156 = call <vilib>:"Std Deviation and Variance.vi"("X"=w306) -> ("mean"=w307:dbl, "standard deviation"=w305:dbl)  [unwired: 1 in, 1 out]
        n157 = call <vilib>:"Std Deviation and Variance.vi"("X"=w298) -> ("mean"=w303:dbl, "standard deviation"=w304:dbl)  [unwired: 1 in, 1 out]
        n158 = call <vilib>:"Std Deviation and Variance.vi"("X"=w294) -> ("mean"=w300:dbl, "standard deviation"=w299:dbl)  [unwired: 1 in, 1 out]
        n159 = call <vilib>:"Std Deviation and Variance.vi"("X"=w296) -> ("mean"=w295:dbl, "standard deviation"=w297:dbl)  [unwired: 1 in, 1 out]
        n160 = call <vilib>:"Std Deviation and Variance.vi"("X"=w319) -> ("mean"=w318:dbl, "standard deviation"=w320:dbl)  [unwired: 1 in, 1 out]
        n161 = call <vilib>:"Std Deviation and Variance.vi"("X"=w316) -> ("mean"=w317:dbl, "standard deviation"=w315:dbl)  [unwired: 1 in, 1 out]
        n162 = call <vilib>:"Std Deviation and Variance.vi"("X"=w313) -> ("mean"=w312:dbl, "standard deviation"=w314:dbl)  [unwired: 1 in, 1 out]
        n163 = call <vilib>:"Std Deviation and Variance.vi"("X"=w290) -> ("mean"=w291:dbl, "standard deviation"=w289:dbl)  [unwired: 1 in, 1 out]
        n164 = call <vilib>:"Std Deviation and Variance.vi"("X"=w287) -> ("mean"=w286:dbl, "standard deviation"=w288:dbl)  [unwired: 1 in, 1 out]
        n165 = call <vilib>:"Std Deviation and Variance.vi"("X"=w282) -> ("mean"=w281:dbl, "standard deviation"=w283:dbl)  [unwired: 1 in, 1 out]
        n166 = call <vilib>:"Std Deviation and Variance.vi"("X"=w279) -> ("mean"=w280:dbl, "standard deviation"=w278:dbl)  [unwired: 1 in, 1 out]
        n167 = Divide(x=w409, y=w410) -> (x/y=w348:dbl)
        n168 = Divide(x=w408, y=w407) -> (x/y=w398:dbl)
        n169 = Divide(x=w405, y=w406) -> (x/y=w397:dbl)
        n170 = Divide(x=w404, y=w403) -> (x/y=w396:dbl)
        n171 = Divide(x=w369, y=w370) -> (x/y=w371:dbl)
        n172 = Divide(x=w324, y=w325) -> (x/y=w326:dbl)
        n173 = Divide(x=w321, y=w322) -> (x/y=w323:dbl)
        n174 = Divide(x=w382, y=w380) -> (x/y=w383:dbl)
        n175 = Divide(x=w378, y=w379) -> (x/y=w377:dbl)
        n176 = Divide(x=w375, y=w374) -> (x/y=w376:dbl)
        n177 = Divide(x=w366, y=w368) -> (x/y=w364:dbl)
        n178 = Divide(x=w393, y=w395) -> (x/y=w386:dbl)
        n179 = Divide(x=w392, y=w390) -> (x/y=w385:dbl)
        n180 = Divide(x=w387, y=w389) -> (x/y=w384:dbl)
        n181 = Divide(x=w362, y=w360) -> (x/y=w363:dbl)
        n182 = Divide(x=w357, y=w359) -> (x/y=w356:dbl)
        n183 = Divide(x=w331, y=w354) -> (x/y=w355:dbl)
        n184 = Divide(x=w307, y=w305) -> (x/y=w308:dbl)
        n185 = Divide(x=w303, y=w304) -> (x/y=w302:dbl)
        n186 = Divide(x=w300, y=w299) -> (x/y=w301:dbl)
        n187 = Divide(x=w295, y=w297) -> (x/y=w293:dbl)
        n188 = Divide(x=w318, y=w320) -> (x/y=w311:dbl)
        n189 = Divide(x=w317, y=w315) -> (x/y=w310:dbl)
        n190 = Divide(x=w312, y=w314) -> (x/y=w309:dbl)
        n191 = Divide(x=w291, y=w289) -> (x/y=w292:dbl)
        n192 = Divide(x=w286, y=w288) -> (x/y=w285:dbl)
        n193 = Divide(x=w281, y=w283) -> (x/y=w284:dbl)
        n194 = Divide(x=w280, y=w278) -> (x/y=w277:dbl)
        n195 = Absolute Value(x=w348) -> (abs(x)=→"1环SNR":dbl)
        n196 = Absolute Value(x=w398) -> (abs(x)=→"2环SNR":dbl)
        n197 = Absolute Value(x=w397) -> (abs(x)=→"3环SNR":dbl)
        n198 = Absolute Value(x=w396) -> (abs(x)=→"4环SNR":dbl)
        n199 = Absolute Value(x=w371) -> (abs(x)=→"5环SNR":dbl)
        n200 = Absolute Value(x=w326) -> (abs(x)=→"6环SNR":dbl)
        n201 = Absolute Value(x=w323) -> (abs(x)=→"7环SNR":dbl)
        n202 = Absolute Value(x=w383) -> (abs(x)=→"1-2":dbl)
        n203 = Absolute Value(x=w377) -> (abs(x)=→"1-3":dbl)
        n204 = Absolute Value(x=w376) -> (abs(x)=→"1-4":dbl)
        n205 = Absolute Value(x=w364) -> (abs(x)=→"1-5":dbl)
        n206 = Absolute Value(x=w386) -> (abs(x)=→"2-3":dbl)
        n207 = Absolute Value(x=w385) -> (abs(x)=→"2-4":dbl)
        n208 = Absolute Value(x=w384) -> (abs(x)=→"2-5":dbl)
        n209 = Absolute Value(x=w363) -> (abs(x)=→"3-4":dbl)
        n210 = Absolute Value(x=w356) -> (abs(x)=→"3-5":dbl)
        n211 = Absolute Value(x=w355) -> (abs(x)=→"4-5":dbl)
        n212 = Absolute Value(x=w308) -> (abs(x)=→"1-6":dbl)
        n213 = Absolute Value(x=w302) -> (abs(x)=→"1-7":dbl)
        n214 = Absolute Value(x=w301) -> (abs(x)=→"2-6":dbl)
        n215 = Absolute Value(x=w293) -> (abs(x)=→"2-7":dbl)
        n216 = Absolute Value(x=w311) -> (abs(x)=→"3-6":dbl)
        n217 = Absolute Value(x=w310) -> (abs(x)=→"3-7":dbl)
        n218 = Absolute Value(x=w309) -> (abs(x)=→"4-6":dbl)
        n219 = Absolute Value(x=w292) -> (abs(x)=→"4-7":dbl)
        n220 = Absolute Value(x=w285) -> (abs(x)=→"5-6":dbl)
        n221 = Absolute Value(x=w284) -> (abs(x)=→"5-7":dbl)
        n222 = Absolute Value(x=w277) -> (abs(x)=→"6-7":dbl)
        n223 = call <vilib>:"Add State(s) to Queue__jki_lib_state_machine.vi"("State(s) in (\"\")"=w242) -> ("States Out"=w243:string)  [unwired: 14 in]
      }
      frame "Data: Cleanup" {
        # "#CSM \"Data: Cleanup\"\nCleanup any data and references, here.\n(this is called automatically, by the Macro: Exit)"
        n224 = Unbundle By Name(w416) -> ("Core.Current VI Reference"=w419:refnum<vi>, "Sample Settings"=w415:T17, "Indicators"=w413:T19)
        n225 = call "CSM - Write Configuration Variable.vim"("Section Name (\"\" as Default)"=w414, "Configuration"=w415) -> ("error out"=w412:errorcluster)  [unwired: 6 in, 1 out]
        n226 = call "CSM - Write Configuration Variable.vim"("Section Name (\"\" as Default)"=w414, "error in (no error)"=w412, "Configuration"=w413) -> ()  [unwired: 5 in, 2 out]
        n227 = Close Reference(reference=w419, error in (no error)=w418) -> (error out=w417:errorcluster)
        n228 = call <vilib>:"Add State(s) to Queue__JKI_lib_State_Machine.vi"("State(s) in (\"\")"=w421) -> ("States Out"=w420:string)  [unwired: 14 in]
      }
      frame "---------- UI ----------" {
        # "#CSM \"Category Seperator\"\nDo not put any code in this frame."
        n229 = call <vilib>:"Add State(s) to Queue__JKI_lib_State_Machine.vi"("State(s) in (\"\")"=w424) -> ("States Out"=w423:string)  [unwired: 14 in]
      }
      frame "UI: Initialize" {
        n230 = Unbundle By Name(w427) -> ("子程序？"=w478:bool, "Indicators.控制.信号采集设备和供电"=w477:tag, "Sample Settings.设备信息.光控设备"=w425:tag, "Indicators.控制.自动停止(周期)"=w476:dbl, "Indicators.控制.自动停止(时间, min)"=w475:dbl, "Indicators.控制.测头类型"=w474:T7, "Sample Settings.等待.等待时"=w468:enum16{"无电无光", "有电无光", "无电有光", "有电有光"}, "Sample Settings.等待.等待方式"=w473:bool, "Sample Settings.等待.每x周期/点等待"=w472:i32, "Sample Settings.等待.等待时间(s)"=w471:dbl, "Indicators.控制.测量波长"=w445:T3[], "Sample Settings.测量.每波长测量次数"=w470:i32, "Indicators.校准.温度校准通道"=w464:T6, "Sample Settings.测量控制.测头拿起"=w444:bool, "Sample Settings.图表相关.文件-时间"=w457:string, "Sample Settings.设备信息.环数"=w450:u8, "Sample Settings.校准.暗电流校准值初值"=w454:dbl[], "Indicators.校准.温度校准值（每度）"=w456:dbl[][])
        n231 = property on="时间-周期" class="WFChart (严格)"("History Data"=waveform(i32)[] [] ("历史数据")) -> ()  [unwired: 2 in, 2 out]
        n232 = property on="时间-周期对照" class="Tbl (严格)"("Value"=string[][] [] ("时间-周期对照")) -> ()  [unwired: 2 in, 2 out]
        n233 = control-ref of="波形查看"() -> (w461:refnum<vi>)
        n234 = Equal?(x=w450, y=u8 7) -> (x = y?=w451:bool)
        n235 = control-ref of="控制台"() -> (w462:refnum<vi>)
        n236 = call <vilib>:"Permute.vi"("k"=u32 2, "n"=w450) -> ("nPk"=w448:dbl)
        n237 = Divide(x=w448, y=2.0) -> (x/y=w446:dbl)
        n238 = Build Array(w462, w461) -> (w460:refnum<vi>[])
        n239 = for {
          tunnel: "7" ("标题包含字符串") -> [w484]
          tunnel: w451 -> [w483]
          tunnel: w460 -> [w482] mode=indexing
          n240 = call "选项卡页面可见.vi"("选项卡可见？"=w483, "标题包含字符串"=w484, "选项卡引用"=w482) -> ()  [unwired: 9 in]
        }
        n241 = Array Subset(array=w454, length=w450) -> (w453:dbl[])  [unwired: 1 in]
        n242 = Array Subset(array=w456, length (row)=w446) -> (w455:dbl[][])  [unwired: 3 in]
        n243 = Not(x=w478) -> (.not. x?=w469:bool)
        n244 = local write "测头拿取"(w444) -> ()
        n245 = local write "等待时"(w468) -> ()
        n246 = local write "测头类型"(w474) -> ()
        n247 = local write "等待方式"(w473) -> ()
        n248 = local write "等待时间(s)"(w471) -> ()
        n249 = local write "校准通道"(w464) -> ()
        n250 = local write "测量波长"(w445) -> ()
        n251 = local write "自动停止(周期)"(w476) -> ()
        n252 = local write "每x周期/点等待"(w472) -> ()
        n253 = local write "每波长测量次数"(w470) -> ()
        n254 = local write "数据文件前缀"(w457) -> ()
        n255 = local write "温度校准值（每度）"(w455) -> ()
        n256 = property on="开始" class="Bool"("DisabledEnum"=T11."Enabled" ("禁用")) -> ()  [unwired: 2 in, 2 out]
        n257 = local write "信号采集设备和供电"(w477) -> ()
        n258 = local write "自动停止(时间, min)"(w475) -> ()
        n259 = local write "光控设备"(w425) -> ()
        n260 = local write "暗电流校准值"(w453) -> ()
        n261 = property on="停止" class="Bool"("Visible"=w469) -> ()  [unwired: 2 in, 2 out]
        n262 = Not(x=w444) -> (.not. x?=w443:bool)
        n263 = property on="6环" class="DigNum (严格)"("Visible"=w451) -> ()  [unwired: 2 in, 2 out]
        n264 = property on="7环" class="DigNum (严格)"("Visible"=w451) -> ()  [unwired: 2 in, 2 out]
        n265 = local write "是否保存"(w443) -> ()
        n266 = local write "测头出光"(w443) -> ()
        n267 = Unbundle By Name(w427) -> ("Indicators.波长差分.X"=w442:T3, "Indicators.波长差分.Y"=w441:T3, "Indicators.波长差分.差分X"=w440:T4, "Indicators.波长差分.差分Y"=w439:T4, "Indicators.波长差分.k"=w438:dbl, "Indicators.波长差分.X2"=w437:T3, "Indicators.波长差分.Y2"=w436:T3, "Indicators.波长差分.差分X2"=w435:T4, "Indicators.波长差分.差分Y2"=w434:T4, "Indicators.波长差分.k2"=w433:dbl, "Indicators.波长差分.X3"=w432:T3, "Indicators.波长差分.Y3"=w431:T3, "Indicators.波长差分.差分X3"=w430:T4, "Indicators.波长差分.差分Y3"=w429:T4, "Indicators.波长差分.k3"=w428:dbl)
        n268 = local write "X"(w442) -> ()
        n269 = local write "Y"(w441) -> ()
        n270 = local write "差分X"(w440) -> ()
        n271 = local write "差分Y"(w439) -> ()
        n272 = local write "k"(w438) -> ()
        n273 = local write "X2"(w437) -> ()
        n274 = local write "Y2"(w436) -> ()
        n275 = local write "差分X2"(w435) -> ()
        n276 = local write "差分Y2"(w434) -> ()
        n277 = local write "k2"(w433) -> ()
        n278 = local write "X3"(w432) -> ()
        n279 = local write "Y3"(w431) -> ()
        n280 = local write "差分X3"(w430) -> ()
        n281 = local write "差分Y3"(w429) -> ()
        n282 = local write "k3"(w428) -> ()
        n283 = in-place {
          in-place-border: w458 -> [w481]
          n284 = in-place-cluster #2(w427) -> ()  [unwired: 1 out]
          n285 = in-place-cluster #2("Sample Settings.CSM.CSM Name"=w481) -> (w426:T20)
        }
        n286 = call <vilib>:"Add State(s) to Queue__JKI_lib_State_Machine.vi"("State(s) in (\"\")"=w480) -> ("States Out"=w479:string)  [unwired: 14 in]
        "程序状态" <- "Ready" ("程序状态")
      }
      frame "UI Initialize Start" {
        n287 = in-place {
          w517 = 1 ("Indicators.图表相关.基准索引")
          n288 = in-place-cluster #3(w485) -> ()  [unwired: 30 out]
          n289 = property on="W单环Aa" class="Ring (严格)"() -> ("Strings []"=w535:string[])  [unwired: 2 in, 2 out]
          n290 = Decimal String To Number(string=w535) -> (number=w507:i32[])  [unwired: 2 in, 1 out]
          n291 = local read "每x周期/点等待"() -> (w515:i32)
          n292 = local read "暗电流校准值"() -> (w508:dbl[])
          n293 = local read "等待时间(s)"() -> (w513:dbl)
          n294 = local read "测头拿取"() -> (w509:bool)
          n295 = local read "是否保存"() -> (w510:bool)
          n296 = local read "测头供电"() -> (w511:bool)
          n297 = local read "测头出光"() -> (w512:bool)
          n298 = local read "等待方式"() -> (w514:bool)
          n299 = local read "温度校准值（每度）"() -> (w518:dbl[][])
          n300 = local read "等待时"() -> (w516:enum16{"无电无光", "有电无光", "无电有光", "有电有光"})
          n301 = local write "A | Ad\n基准周期"(w517) -> ()
          n302 = local read "X"() -> (w520:T3)
          n303 = local read "Y"() -> (w521:T3)
          n304 = local read "差分X"() -> (w522:T4)
          n305 = local read "差分Y"() -> (w523:T4)
          n306 = local read "k"() -> (w524:dbl)
          n307 = local read "X2"() -> (w525:T3)
          n308 = local read "Y2"() -> (w526:T3)
          n309 = local read "差分X2"() -> (w527:T4)
          n310 = local read "差分Y2"() -> (w528:T4)
          n311 = local read "k2"() -> (w529:dbl)
          n312 = local read "X3"() -> (w530:T3)
          n313 = local read "Y3"() -> (w531:T3)
          n314 = local read "差分X3"() -> (w532:T4)
          n315 = local read "差分Y3"() -> (w533:T4)
          n316 = local read "k3"() -> (w534:dbl)
          n317 = in-place-cluster #3("Sample Settings.设备信息.光谱保存路径"=path "D:/sunrise/data" ("存储路径"), "Sample Settings.测量.每波长测量次数"="每波长测量次数", "Sample Settings.测量.波长"=w507, "Sample Settings.校准.暗电流校准值初值"=w508, "Sample Settings.测量控制.测头拿起"=w509, "Sample Settings.测量控制.起始保存"=w510, "Sample Settings.测量控制.测头供电"=w511, "Sample Settings.测量控制.测头出光"=w512, "Sample Settings.等待.等待时间(s)"=w513, "Sample Settings.等待.等待方式"=w514, "Sample Settings.等待.每x周期/点等待"=w515, "Sample Settings.等待.等待时"=w516, "Sample Settings.设备信息.光控设备"="光控设备", "Indicators.图表相关.基准索引"=w517, "Indicators.校准.温度校准值（每度）"=w518, "Indicators.波长差分.X"=w520, "Indicators.波长差分.Y"=w521, "Indicators.波长差分.差分X"=w522, "Indicators.波长差分.差分Y"=w523, "Indicators.波长差分.k"=w524, "Indicators.波长差分.X2"=w525, "Indicators.波长差分.Y2"=w526, "Indicators.波长差分.差分X2"=w527, "Indicators.波长差分.差分Y2"=w528, "Indicators.波长差分.k2"=w529, "Indicators.波长差分.X3"=w530, "Indicators.波长差分.Y3"=w531, "Indicators.波长差分.差分X3"=w532, "Indicators.波长差分.差分Y3"=w533, "Indicators.波长差分.k3"=w534) -> (w486:T20)
        }
        n318 = Unbundle By Name(w485) -> ("Sample Settings.设备信息.环数"=w497:u8)
        n319 = control-ref of="波形查看"() -> (w502:refnum<vi>)
        n320 = Equal?(x=w497, y=u8 7) -> (x = y?=w489:bool)
        n321 = control-ref of="控制台"() -> (w503:refnum<vi>)
        n322 = local read "计时方式"() -> (w487:bool)
        n323 = Build Array(w503, w502) -> (w501:refnum<vi>[])
        n324 = case shown="True" w487 {
          frame False {
          }
          frame True {
            n325 = local write "开始/清零"(TRUE ("暂停/继续")) -> ()
          }
        }
        n326 = for {
          tunnel: "7" ("标题包含字符串") -> [w539]
          tunnel: w489 -> [w538]
          tunnel: w501 -> [w537] mode=indexing
          n327 = call "选项卡页面可见.vi"("选项卡可见？"=w538, "标题包含字符串"=w539, "选项卡引用"=w537) -> ()  [unwired: 9 in]
        }
        n328 = local write "程序状态"("开始" ("程序状态")) -> ()
        n329 = property on="开始" class="Bool"("DisabledEnum"=T11."Disabled and Grayed Out" ("禁用")) -> ()  [unwired: 2 in, 2 out]
        n330 = property on="6环" class="DigNum (严格)"("Visible"=w489) -> ()  [unwired: 2 in, 2 out]
        n331 = property on="7环" class="DigNum (严格)"("Visible"=w489) -> ()  [unwired: 2 in, 2 out]
        n332 = Unbundle By Name(w486) -> ("Sample Settings"=w495:T17)
        n333 = call "Convert Data To API String Arguments.vim"("Data"=w495) -> ("API String"=w496:string)  [unwired: 7 in, 1 out]
        n334 = call-poly <userlib>:"Build Message with Arguments++.vi"("States With Replace Token"="API: Start >> <param> -@ Acquisition - <1>\nAPI: Start >> <param> -@ Logging - <1>" ("State"), "<param>"=w496, "<1>"=w490) -> ("States"=w492:string)  [unwired: 12 in]
        n335 = call <vilib>:"Add State(s) to Queue__jki_lib_state_machine.vi"("State(s) in Front (\"\")"=w492, "State(s) in (\"\")"=w493) -> ("States Out"=w494:string)  [unwired: 13 in]
      }
      frame "UI: Update Graph" {
        n336 = Unbundle By Name(w560) -> ("Time and Data.当前运行信息.当前周期"=w549:i32, "Indicators.图表相关.程序开始时间"=w548:timestamp, "Sample Settings.测量控制.测头拿起"=w550:bool, "Sample Settings.设备信息.环数"=w553:u8, "Time and Data.Logging Settings.周期结束？"=w546:bool, "Time and Data.Logging Settings.波长结束？"=w540:bool, "Time and Data.采集时间"=w547:timestamp)
        n337 = case shown="True" w546 {
          tunnel: w549 -> [_ w574]
          tunnel: w547 -> [_ w573]
          frame False {
          }
          frame True {
            n338 = Format Date/Time String(time format string (%c)="%H: %M: %S" ("时间格式字符串(%c)"), seconds (now)=w573) -> (date/time string=w578:string)  [unwired: 1 in]
            n339 = Number To Decimal String(number=w574) -> (decimal integer string=w580:string)  [unwired: 1 in]
            n340 = Build Array(w580, w578) -> (w577:string[])
            n341 = Build Array(w574) -> (w583:i32[])
            n342 = feedback #4(string[][] []) -> (w576:string[][])
            n343 = Build Array (concatenate)(w576, w577) -> (w581:string[][])
            "时间-周期对照" <- w581
            n344 = feedback-in #4(w581) -> ()
            n345 = Bundle By Name("Y"=w583, "t0"=w573) -> (→"时间-周期":waveform(i32))  [unwired: 1 in]
          }
        }
        n346 = Get Date/Time In Seconds() -> (seconds since 1Jan1904=w566:timestamp)
        n347 = Subtract(x=w566, y=w548) -> (x-y=w565:dbl)
        n348 = Equal?(x=w553, y=u8 7) -> (x = y?=w545:bool)
        n349 = Divide(x=w565, y=60.0) -> (x/y=w562:dbl)
        "已运行时间(min)" <- w562
        n350 = Greater?(x=w562, y="自动停止(时间, min)") -> (0:w563:bool)
        n351 = Greater?(x=w549, y="自动停止(周期)") -> (0:w567:bool)
        n352 = Compound Arithmetic op=OR ("复合运算")(w567, w563) -> (w558:bool)
        n353 = case shown="True" w546 {
          tunnel: ["" ("State(s) at Back (\"\")") "UI: Update Graph_Diff_Wave" ("State(s) at Back (\"\")")] -> w554
          frame False {
          }
          frame True {
          }
        }
        n354 = case shown="True" w540 {
          tunnel: ["" ("State(s) at Back (\"\")") "Data: Update SNR" ("State(s) in (\"\")")] -> w541
          frame False {
          }
          frame True {
          }
        }
        n355 = case shown="True" w545 {
          tunnel: ["" ("State(s) in (\"\")") "UI: Update Graph_Diff_7R" ("State(s) in (\"\")")] -> w555
          frame False {
          }
          frame True {
          }
        }
        n356 = call <vilib>:"Add State(s) to Queue__JKI_lib_State_Machine.vi"("State(s) in Front (\"\")"="UI: Update Graph_Single\nUI: Update Graph_Diff\n\nUI: Update Graph_Single_LT\nUI: Update Graph_Diff_LT1\nUI: Update Graph_Diff_LT2\nUI: Update Graph_Diff_LT3\n" ("f"), "State(s) in (\"\")"=w555, "State(s) at Back (\"\")"=w554) -> ("States Out"=w542:string)  [unwired: 12 in]
        n357 = call <vilib>:"Add State(s) to Queue__jki_lib_state_machine.vi"("State(s) in (\"\")"=w542, "State(s) at Back (\"\")"=w541) -> ("States Out"=w543:string)  [unwired: 13 in]
        n358 = Select(t="", s=w550, f=w543) -> (s? t:f=w552:string)
        n359 = Select(t="Macro: Exit" ("State(s) in Front (\"\")"), s=w558, f=w552) -> (s? t:f=w557:string)
        n360 = call <vilib>:"Add State(s) to Queue__JKI_lib_State_Machine.vi"("State(s) in Front (\"\")"=w557, "State(s) in (\"\")"=w570) -> ("States Out"=w569:string)  [unwired: 13 in]
      }
      frame "UI: Update Graph_Single" {
        # "短期-单环"
        n361 = Unbundle By Name(w597) -> ("Time and Data.当前运行信息.当前索引子集"=w589:i8[], "Time and Data.Data"=w598:dbl[])
        n362 = Index Array(array=w589) -> (element=w588:i8)  [unwired: 1 in]
        n363 = Index Array(array=w598) -> (element #1=w596:dbl, element #2=w595:dbl, element #3=w594:dbl, element #4=w593:dbl, element #5=w592:dbl, element #6=w591:dbl, element #7=w590:dbl)  [unwired: 7 in]
        n364 = case shown="1" w588 {
          tunnel: w596 -> [_ w709 w714 w717 w720 w723 w726]
          frame -1, Default {
          }
          frame 0 {
            n365 = call "信号收集器2"("Signals"=w709) -> ("Collected Signals"=w711:dynamicdata)  [unwired: 9 in, 1 out]
            n366 = call "从动态数据转换5"("Dynamic Data Type"=w711) -> ("Array"=→"1050":dbl[])  [unwired: 3 in]
          }
          frame 1 {
            n367 = call "信号收集器"("Signals"=w714) -> ("Collected Signals"=w712:dynamicdata)  [unwired: 9 in, 1 out]
            n368 = call "从动态数据转换6"("Dynamic Data Type"=w712) -> ("Array"=→"1213":dbl[])  [unwired: 3 in]
          }
          frame 2 {
            n369 = call "信号收集器3"("Signals"=w717) -> ("Collected Signals"=w715:dynamicdata)  [unwired: 9 in, 1 out]
            n370 = call "从动态数据转换7"("Dynamic Data Type"=w715) -> ("Array"=→"1314":dbl[])  [unwired: 3 in]
          }
          frame 3 {
            n371 = call "信号收集器4"("Signals"=w720) -> ("Collected Signals"=w719:dynamicdata)  [unwired: 9 in, 1 out]
            n372 = call "从动态数据转换8"("Dynamic Data Type"=w719) -> ("Array"=→"1409":dbl[])  [unwired: 3 in]
          }
          frame 4 {
            n373 = call "信号收集器5"("Signals"=w723) -> ("Collected Signals"=w721:dynamicdata)  [unwired: 9 in, 1 out]
            n374 = call "从动态数据转换9"("Dynamic Data Type"=w721) -> ("Array"=→"1550":dbl[])  [unwired: 3 in]
          }
          frame 5 {
            n375 = call "信号收集器6"("Signals"=w726) -> ("Collected Signals"=w725:dynamicdata)  [unwired: 9 in, 1 out]
            n376 = call "从动态数据转换11"("Dynamic Data Type"=w725) -> ("Array"=→"1609":dbl[])  [unwired: 3 in]
          }
        }
        n377 = case shown="2" w588 {
          tunnel: w595 -> [_ w693 w696 w699 w702 w705 w708]
          frame -1, Default {
          }
          frame 0 {
            n378 = call "信号收集器7"("Signals"=w693) -> ("Collected Signals"=w692:dynamicdata)  [unwired: 9 in, 1 out]
            n379 = call "从动态数据转换12"("Dynamic Data Type"=w692) -> ("Array"=→"1050 2":dbl[])  [unwired: 3 in]
          }
          frame 1 {
            n380 = call "信号收集器8"("Signals"=w696) -> ("Collected Signals"=w695:dynamicdata)  [unwired: 9 in, 1 out]
            n381 = call "从动态数据转换13"("Dynamic Data Type"=w695) -> ("Array"=→"1213 3":dbl[])  [unwired: 3 in]
          }
          frame 2 {
            n382 = call "信号收集器9"("Signals"=w699) -> ("Collected Signals"=w697:dynamicdata)  [unwired: 9 in, 1 out]
            n383 = call "从动态数据转换14"("Dynamic Data Type"=w697) -> ("Array"=→"1314 2":dbl[])  [unwired: 3 in]
          }
          frame 3 {
            n384 = call "信号收集器10"("Signals"=w702) -> ("Collected Signals"=w700:dynamicdata)  [unwired: 9 in, 1 out]
            n385 = call "从动态数据转换16"("Dynamic Data Type"=w700) -> ("Array"=→"1409 3":dbl[])  [unwired: 3 in]
          }
          frame 4 {
            n386 = call "信号收集器11"("Signals"=w705) -> ("Collected Signals"=w703:dynamicdata)  [unwired: 9 in, 1 out]
            n387 = call "从动态数据转换17"("Dynamic Data Type"=w703) -> ("Array"=→"1550 3":dbl[])  [unwired: 3 in]
          }
          frame 5 {
            n388 = call "信号收集器12"("Signals"=w708) -> ("Collected Signals"=w707:dynamicdata)  [unwired: 9 in, 1 out]
            n389 = call "从动态数据转换10"("Dynamic Data Type"=w707) -> ("Array"=→"1609 3":dbl[])  [unwired: 3 in]
          }
        }
        n390 = case shown="4" w588 {
          tunnel: w593 -> [_ w655 w660 w663 w666 w667 w672]
          frame -1, Default {
          }
          frame 0 {
            n391 = call "信号收集器25"("Signals"=w655) -> ("Collected Signals"=w656:dynamicdata)  [unwired: 9 in, 1 out]
            n392 = call "从动态数据转换30"("Dynamic Data Type"=w656) -> ("Array"=→"1050 4":dbl[])  [unwired: 3 in]
          }
          frame 1 {
            n393 = call "信号收集器26"("Signals"=w660) -> ("Collected Signals"=w659:dynamicdata)  [unwired: 9 in, 1 out]
            n394 = call "从动态数据转换31"("Dynamic Data Type"=w659) -> ("Array"=→"1213 4":dbl[])  [unwired: 3 in]
          }
          frame 2 {
            n395 = call "信号收集器27"("Signals"=w663) -> ("Collected Signals"=w661:dynamicdata)  [unwired: 9 in, 1 out]
            n396 = call "从动态数据转换32"("Dynamic Data Type"=w661) -> ("Array"=→"1314 4":dbl[])  [unwired: 3 in]
          }
          frame 3 {
            n397 = call "信号收集器28"("Signals"=w666) -> ("Collected Signals"=w664:dynamicdata)  [unwired: 9 in, 1 out]
            n398 = call "从动态数据转换33"("Dynamic Data Type"=w664) -> ("Array"=→"1409 4":dbl[])  [unwired: 3 in]
          }
          frame 4 {
            n399 = call "信号收集器29"("Signals"=w667) -> ("Collected Signals"=w668:dynamicdata)  [unwired: 9 in, 1 out]
            n400 = call "从动态数据转换34"("Dynamic Data Type"=w668) -> ("Array"=→"1550 4":dbl[])  [unwired: 3 in]
          }
          frame 5 {
            n401 = call "信号收集器30"("Signals"=w672) -> ("Collected Signals"=w670:dynamicdata)  [unwired: 9 in, 1 out]
            n402 = call "从动态数据转换19"("Dynamic Data Type"=w670) -> ("Array"=→"1609 4":dbl[])  [unwired: 3 in]
          }
        }
        n403 = case shown="3" w588 {
          tunnel: w590 -> [_ w602 w606 w609 w612 w614 w618]
          frame -1, Default {
          }
          frame 0 {
            n404 = call "信号收集器97"("Signals"=w602) -> ("Collected Signals"=w603:dynamicdata)  [unwired: 9 in, 1 out]
            n405 = call "从动态数据转换97"("Dynamic Data Type"=w603) -> ("Array"=→"1050 16":dbl[])  [unwired: 3 in]
          }
          frame 1 {
            n406 = call "信号收集器98"("Signals"=w606) -> ("Collected Signals"=w605:dynamicdata)  [unwired: 9 in, 1 out]
            n407 = call "从动态数据转换98"("Dynamic Data Type"=w605) -> ("Array"=→"1213 16":dbl[])  [unwired: 3 in]
          }
          frame 2 {
            n408 = call "信号收集器99"("Signals"=w609) -> ("Collected Signals"=w608:dynamicdata)  [unwired: 9 in, 1 out]
            n409 = call "从动态数据转换99"("Dynamic Data Type"=w608) -> ("Array"=→"1314 16":dbl[])  [unwired: 3 in]
          }
          frame 3 {
            n410 = call "信号收集器100"("Signals"=w612) -> ("Collected Signals"=w611:dynamicdata)  [unwired: 9 in, 1 out]
            n411 = call "从动态数据转换100"("Dynamic Data Type"=w611) -> ("Array"=→"1409 16":dbl[])  [unwired: 3 in]
          }
          frame 4 {
            n412 = call "信号收集器101"("Signals"=w614) -> ("Collected Signals"=w615:dynamicdata)  [unwired: 9 in, 1 out]
            n413 = call "从动态数据转换101"("Dynamic Data Type"=w615) -> ("Array"=→"1550 14":dbl[])  [unwired: 3 in]
          }
          frame 5 {
            n414 = call "信号收集器102"("Signals"=w618) -> ("Collected Signals"=w617:dynamicdata)  [unwired: 9 in, 1 out]
            n415 = call "从动态数据转换102"("Dynamic Data Type"=w617) -> ("Array"=→"1609 16":dbl[])  [unwired: 3 in]
          }
        }
        n416 = case shown="3" w588 {
          tunnel: w591 -> [_ w620 w624 w627 w630 w632 w636]
          frame -1, Default {
          }
          frame 0 {
            n417 = call "信号收集器91"("Signals"=w620) -> ("Collected Signals"=w621:dynamicdata)  [unwired: 9 in, 1 out]
            n418 = call "从动态数据转换"("Dynamic Data Type"=w621) -> ("Array"=→"1050 15":dbl[])  [unwired: 3 in]
          }
          frame 1 {
            n419 = call "信号收集器92"("Signals"=w624) -> ("Collected Signals"=w623:dynamicdata)  [unwired: 9 in, 1 out]
            n420 = call "从动态数据转换2"("Dynamic Data Type"=w623) -> ("Array"=→"1213 15":dbl[])  [unwired: 3 in]
          }
          frame 2 {
            n421 = call "信号收集器93"("Signals"=w627) -> ("Collected Signals"=w626:dynamicdata)  [unwired: 9 in, 1 out]
            n422 = call "从动态数据转换3"("Dynamic Data Type"=w626) -> ("Array"=→"1314 15":dbl[])  [unwired: 3 in]
          }
          frame 3 {
            n423 = call "信号收集器94"("Signals"=w630) -> ("Collected Signals"=w629:dynamicdata)  [unwired: 9 in, 1 out]
            n424 = call "从动态数据转换4"("Dynamic Data Type"=w629) -> ("Array"=→"1409 15":dbl[])  [unwired: 3 in]
          }
          frame 4 {
            n425 = call "信号收集器95"("Signals"=w632) -> ("Collected Signals"=w633:dynamicdata)  [unwired: 9 in, 1 out]
            n426 = call "从动态数据转换95"("Dynamic Data Type"=w633) -> ("Array"=→"1550 9":dbl[])  [unwired: 3 in]
          }
          frame 5 {
            n427 = call "信号收集器96"("Signals"=w636) -> ("Collected Signals"=w635:dynamicdata)  [unwired: 9 in, 1 out]
            n428 = call "从动态数据转换96"("Dynamic Data Type"=w635) -> ("Array"=→"1609 15":dbl[])  [unwired: 3 in]
          }
        }
        n429 = case shown="3" w588 {
          tunnel: w594 -> [_ w673 w678 w681 w684 w685 w690]
          frame -1, Default {
          }
          frame 0 {
            n430 = call "信号收集器19"("Signals"=w673) -> ("Collected Signals"=w674:dynamicdata)  [unwired: 9 in, 1 out]
            n431 = call "从动态数据转换18"("Dynamic Data Type"=w674) -> ("Array"=→"1050 5":dbl[])  [unwired: 3 in]
          }
          frame 1 {
            n432 = call "信号收集器20"("Signals"=w678) -> ("Collected Signals"=w676:dynamicdata)  [unwired: 9 in, 1 out]
            n433 = call "从动态数据转换25"("Dynamic Data Type"=w676) -> ("Array"=→"1213 5":dbl[])  [unwired: 3 in]
          }
          frame 2 {
            n434 = call "信号收集器21"("Signals"=w681) -> ("Collected Signals"=w679:dynamicdata)  [unwired: 9 in, 1 out]
            n435 = call "从动态数据转换26"("Dynamic Data Type"=w679) -> ("Array"=→"1314 5":dbl[])  [unwired: 3 in]
          }
          frame 3 {
            n436 = call "信号收集器22"("Signals"=w684) -> ("Collected Signals"=w682:dynamicdata)  [unwired: 9 in, 1 out]
            n437 = call "从动态数据转换27"("Dynamic Data Type"=w682) -> ("Array"=→"1409 5":dbl[])  [unwired: 3 in]
          }
          frame 4 {
            n438 = call "信号收集器23"("Signals"=w685) -> ("Collected Signals"=w686:dynamicdata)  [unwired: 9 in, 1 out]
            n439 = call "从动态数据转换28"("Dynamic Data Type"=w686) -> ("Array"=→"1550 5":dbl[])  [unwired: 3 in]
          }
          frame 5 {
            n440 = call "信号收集器24"("Signals"=w690) -> ("Collected Signals"=w688:dynamicdata)  [unwired: 9 in, 1 out]
            n441 = call "从动态数据转换29"("Dynamic Data Type"=w688) -> ("Array"=→"1609 5":dbl[])  [unwired: 3 in]
          }
        }
        n442 = case shown="0" w588 {
          tunnel: w592 -> [_ w637 w642 w645 w648 w649 w654]
          frame -1, Default {
          }
          frame 0 {
            n443 = call "信号收集器31"("Signals"=w637) -> ("Collected Signals"=w638:dynamicdata)  [unwired: 9 in, 1 out]
            n444 = call "从动态数据转换36"("Dynamic Data Type"=w638) -> ("Array"=→"1050 3":dbl[])  [unwired: 3 in]
          }
          frame 1 {
            n445 = call "信号收集器32"("Signals"=w642) -> ("Collected Signals"=w640:dynamicdata)  [unwired: 9 in, 1 out]
            n446 = call "从动态数据转换37"("Dynamic Data Type"=w640) -> ("Array"=→"1213 2":dbl[])  [unwired: 3 in]
          }
          frame 2 {
            n447 = call "信号收集器33"("Signals"=w645) -> ("Collected Signals"=w643:dynamicdata)  [unwired: 9 in, 1 out]
            n448 = call "从动态数据转换38"("Dynamic Data Type"=w643) -> ("Array"=→"1314 3":dbl[])  [unwired: 3 in]
          }
          frame 3 {
            n449 = call "信号收集器34"("Signals"=w648) -> ("Collected Signals"=w646:dynamicdata)  [unwired: 9 in, 1 out]
            n450 = call "从动态数据转换39"("Dynamic Data Type"=w646) -> ("Array"=→"1409 2":dbl[])  [unwired: 3 in]
          }
          frame 4 {
            n451 = call "信号收集器35"("Signals"=w649) -> ("Collected Signals"=w650:dynamicdata)  [unwired: 9 in, 1 out]
            n452 = call "从动态数据转换40"("Dynamic Data Type"=w650) -> ("Array"=→"1550 2":dbl[])  [unwired: 3 in]
          }
          frame 5 {
            n453 = call "信号收集器36"("Signals"=w654) -> ("Collected Signals"=w653:dynamicdata)  [unwired: 9 in, 1 out]
            n454 = call "从动态数据转换35"("Dynamic Data Type"=w653) -> ("Array"=→"1609 2":dbl[])  [unwired: 3 in]
          }
        }
        n455 = call <vilib>:"Add State(s) to Queue__JKI_lib_State_Machine.vi"("State(s) in (\"\")"=w600) -> ("States Out"=w599:string)  [unwired: 14 in]
      }
      frame "UI: Update Graph_Diff" {
        # "短期-差分（五环）"
        # "2-5"
        # "3-5"
        # "2-4"
        # "4-5"
        # "3-4"
        # "2-3"
        # "1-5"
        # "1-4"
        # "1-3"
        # "1-2"
        n456 = Unbundle By Name(w735) -> ("Time and Data.当前运行信息.当前索引子集"=w729:i8[], "Time and Data.Data"=w736:dbl[], "Sample Settings.校准.温度校准值"=w728:dbl[])
        n457 = Index Array(array=w729) -> (element=w727:i8)  [unwired: 1 in]
        n458 = Index Array(array=w736) -> (element #1=w734:dbl, element #2=w733:dbl, element #3=w732:dbl, element #4=w731:dbl, element #5=w730:dbl)  [unwired: 7 in, 2 out]
        n459 = xnode "公式25"("X1"=w733, "X2"=w730) -> ("结果"=w757:dbl)  [unwired: 1 in, 1 out]
        n460 = xnode "公式34"("X1"=w732, "X2"=w731) -> ("结果"=w754:dbl)  [unwired: 1 in, 1 out]
        n461 = xnode "公式35"("X1"=w732, "X2"=w730) -> ("结果"=w751:dbl)  [unwired: 1 in, 1 out]
        n462 = xnode "公式45"("X1"=w731, "X2"=w730) -> ("结果"=w748:dbl)  [unwired: 1 in, 1 out]
        n463 = xnode "公式12"("X1"=w734, "X2"=w733) -> ("结果"=w775:dbl)  [unwired: 1 in, 1 out]
        n464 = xnode "公式13"("X1"=w734, "X2"=w732) -> ("结果"=w772:dbl)  [unwired: 1 in, 1 out]
        n465 = xnode "公式14"("X1"=w734, "X2"=w731) -> ("结果"=w769:dbl)  [unwired: 1 in, 1 out]
        n466 = xnode "公式15"("X1"=w734, "X2"=w730) -> ("结果"=w763:dbl)  [unwired: 1 in, 1 out]
        n467 = xnode "公式23"("X1"=w733, "X2"=w732) -> ("结果"=w765:dbl)  [unwired: 1 in, 1 out]
        n468 = xnode "公式24"("X1"=w733, "X2"=w731) -> ("结果"=w759:dbl)  [unwired: 1 in, 1 out]
        n469 = Index Array(array=w728, index=9 ("索引")) -> (element=w749:dbl)
        n470 = Index Array(array=w728, index=0 ("索引")) -> (element=w776:dbl)
        n471 = Index Array(array=w728, index=7 ("索引")) -> (element=w755:dbl)
        n472 = Index Array(array=w728, index=8 ("索引")) -> (element=w752:dbl)
        n473 = Index Array(array=w728, index=1 ("索引")) -> (element=w773:dbl)
        n474 = Index Array(array=w728, index=3 ("索引")) -> (element=w766:dbl)
        n475 = Index Array(array=w728, index=4 ("索引")) -> (element=w767:dbl)
        n476 = Index Array(array=w728, index=2 ("索引")) -> (element=w770:dbl)
        n477 = Index Array(array=w728, index=6 ("索引")) -> (element=w760:dbl)
        n478 = Index Array(array=w728, index=5 ("索引")) -> (element=w761:dbl)
        n479 = Subtract(x=w748, y=w749) -> (x-y=w747:dbl)
        n480 = Subtract(x=w775, y=w776) -> (x-y=w774:dbl)
        n481 = Subtract(x=w754, y=w755) -> (x-y=w753:dbl)
        n482 = Subtract(x=w751, y=w752) -> (x-y=w750:dbl)
        n483 = Subtract(x=w772, y=w773) -> (x-y=w771:dbl)
        n484 = Subtract(x=w763, y=w766) -> (x-y=w762:dbl)
        n485 = Subtract(x=w765, y=w767) -> (x-y=w764:dbl)
        n486 = Subtract(x=w769, y=w770) -> (x-y=w768:dbl)
        n487 = Subtract(x=w757, y=w760) -> (x-y=w756:dbl)
        n488 = Subtract(x=w759, y=w761) -> (x-y=w758:dbl)
        n489 = case shown="3" w727 {
          tunnel: w774 -> [_ w941 w946 w949 w952 w953 w958]
          frame -1, Default {
          }
          frame 0 {
            n490 = call "信号收集器13"("Signals"=w941) -> ("Collected Signals"=w943:dynamicdata)  [unwired: 9 in, 1 out]
            n491 = call "从动态数据转换24"("Dynamic Data Type"=w943) -> ("Array"=→"1050":dbl[])  [unwired: 3 in]
          }
          frame 1 {
            n492 = call "信号收集器14"("Signals"=w946) -> ("Collected Signals"=w944:dynamicdata)  [unwired: 9 in, 1 out]
            n493 = call "从动态数据转换15"("Dynamic Data Type"=w944) -> ("Array"=→"1213":dbl[])  [unwired: 3 in]
          }
          frame 2 {
            n494 = call "信号收集器15"("Signals"=w949) -> ("Collected Signals"=w948:dynamicdata)  [unwired: 9 in, 1 out]
            n495 = call "从动态数据转换20"("Dynamic Data Type"=w948) -> ("Array"=→"1314":dbl[])  [unwired: 3 in]
          }
          frame 3 {
            n496 = call "信号收集器16"("Signals"=w952) -> ("Collected Signals"=w951:dynamicdata)  [unwired: 9 in, 1 out]
            n497 = call "从动态数据转换21"("Dynamic Data Type"=w951) -> ("Array"=→"1409":dbl[])  [unwired: 3 in]
          }
          frame 4 {
            n498 = call "信号收集器17"("Signals"=w953) -> ("Collected Signals"=w954:dynamicdata)  [unwired: 9 in, 1 out]
            n499 = call "从动态数据转换22"("Dynamic Data Type"=w954) -> ("Array"=→"1550":dbl[])  [unwired: 3 in]
          }
          frame 5 {
            n500 = call "信号收集器18"("Signals"=w958) -> ("Collected Signals"=w957:dynamicdata)  [unwired: 9 in, 1 out]
            n501 = call "从动态数据转换23"("Dynamic Data Type"=w957) -> ("Array"=→"1609":dbl[])  [unwired: 3 in]
          }
        }
        n502 = case shown="0" w727 {
          tunnel: w753 -> [_ w851 w856 w859 w862 w863 w866]
          frame -1, Default {
          }
          frame 0 {
            n503 = call "信号收集器61"("Signals"=w851) -> ("Collected Signals"=w853:dynamicdata)  [unwired: 9 in, 1 out]
            n504 = call "从动态数据转换67"("Dynamic Data Type"=w853) -> ("Array"=→"1050 10":dbl[])  [unwired: 3 in]
          }
          frame 1 {
            n505 = call "信号收集器62"("Signals"=w856) -> ("Collected Signals"=w855:dynamicdata)  [unwired: 9 in, 1 out]
            n506 = call "从动态数据转换68"("Dynamic Data Type"=w855) -> ("Array"=→"1213 10":dbl[])  [unwired: 3 in]
          }
          frame 2 {
            n507 = call "信号收集器63"("Signals"=w859) -> ("Collected Signals"=w858:dynamicdata)  [unwired: 9 in, 1 out]
            n508 = call "从动态数据转换69"("Dynamic Data Type"=w858) -> ("Array"=→"1314 10":dbl[])  [unwired: 3 in]
          }
          frame 3 {
            n509 = call "信号收集器64"("Signals"=w862) -> ("Collected Signals"=w861:dynamicdata)  [unwired: 9 in, 1 out]
            n510 = call "从动态数据转换70"("Dynamic Data Type"=w861) -> ("Array"=→"1409 10":dbl[])  [unwired: 3 in]
          }
          frame 4 {
            n511 = call "信号收集器65"("Signals"=w863) -> ("Collected Signals"=w865:dynamicdata)  [unwired: 9 in, 1 out]
            n512 = call "从动态数据转换65"("Dynamic Data Type"=w865) -> ("Array"=→"1550 10":dbl[])  [unwired: 3 in]
          }
          frame 5 {
            n513 = call "信号收集器66"("Signals"=w866) -> ("Collected Signals"=w868:dynamicdata)  [unwired: 9 in, 1 out]
            n514 = call "从动态数据转换66"("Dynamic Data Type"=w868) -> ("Array"=→"1609 10":dbl[])  [unwired: 3 in]
          }
        }
        n515 = case shown="5" w727 {
          tunnel: w750 -> [_ w797 w802 w805 w808 w809 w814]
          frame -1, Default {
          }
          frame 0 {
            n516 = call "信号收集器79"("Signals"=w797) -> ("Collected Signals"=w798:dynamicdata)  [unwired: 9 in, 1 out]
            n517 = call "从动态数据转换89"("Dynamic Data Type"=w798) -> ("Array"=→"1050 13":dbl[])  [unwired: 3 in]
          }
          frame 1 {
            n518 = call "信号收集器80"("Signals"=w802) -> ("Collected Signals"=w801:dynamicdata)  [unwired: 9 in, 1 out]
            n519 = call "从动态数据转换88"("Dynamic Data Type"=w801) -> ("Array"=→"1213 13":dbl[])  [unwired: 3 in]
          }
          frame 2 {
            n520 = call "信号收集器81"("Signals"=w805) -> ("Collected Signals"=w803:dynamicdata)  [unwired: 9 in, 1 out]
            n521 = call "从动态数据转换83"("Dynamic Data Type"=w803) -> ("Array"=→"1314 13":dbl[])  [unwired: 3 in]
          }
          frame 3 {
            n522 = call "信号收集器82"("Signals"=w808) -> ("Collected Signals"=w807:dynamicdata)  [unwired: 9 in, 1 out]
            n523 = call "从动态数据转换84"("Dynamic Data Type"=w807) -> ("Array"=→"1409 13":dbl[])  [unwired: 3 in]
          }
          frame 4 {
            n524 = call "信号收集器83"("Signals"=w809) -> ("Collected Signals"=w810:dynamicdata)  [unwired: 9 in, 1 out]
            n525 = call "从动态数据转换85"("Dynamic Data Type"=w810) -> ("Array"=→"1550 13":dbl[])  [unwired: 3 in]
          }
          frame 5 {
            n526 = call "信号收集器84"("Signals"=w814) -> ("Collected Signals"=w813:dynamicdata)  [unwired: 9 in, 1 out]
            n527 = call "从动态数据转换86"("Dynamic Data Type"=w813) -> ("Array"=→"1609 13":dbl[])  [unwired: 3 in]
          }
        }
        n528 = case shown="3" w727 {
          tunnel: w768 -> [_ w905 w910 w913 w916 w917 w922]
          frame -1, Default {
          }
          frame 0 {
            n529 = call "信号收集器43"("Signals"=w905) -> ("Collected Signals"=w907:dynamicdata)  [unwired: 9 in, 1 out]
            n530 = call "从动态数据转换48"("Dynamic Data Type"=w907) -> ("Array"=→"1050 7":dbl[])  [unwired: 3 in]
          }
          frame 1 {
            n531 = call "信号收集器44"("Signals"=w910) -> ("Collected Signals"=w909:dynamicdata)  [unwired: 9 in, 1 out]
            n532 = call "从动态数据转换49"("Dynamic Data Type"=w909) -> ("Array"=→"1213 7":dbl[])  [unwired: 3 in]
          }
          frame 2 {
            n533 = call "信号收集器45"("Signals"=w913) -> ("Collected Signals"=w912:dynamicdata)  [unwired: 9 in, 1 out]
            n534 = call "从动态数据转换50"("Dynamic Data Type"=w912) -> ("Array"=→"1314 7":dbl[])  [unwired: 3 in]
          }
          frame 3 {
            n535 = call "信号收集器46"("Signals"=w916) -> ("Collected Signals"=w915:dynamicdata)  [unwired: 9 in, 1 out]
            n536 = call "从动态数据转换51"("Dynamic Data Type"=w915) -> ("Array"=→"1409 7":dbl[])  [unwired: 3 in]
          }
          frame 4 {
            n537 = call "信号收集器47"("Signals"=w917) -> ("Collected Signals"=w919:dynamicdata)  [unwired: 9 in, 1 out]
            n538 = call "从动态数据转换52"("Dynamic Data Type"=w919) -> ("Array"=→"1550 7":dbl[])  [unwired: 3 in]
          }
          frame 5 {
            n539 = call "信号收集器48"("Signals"=w922) -> ("Collected Signals"=w921:dynamicdata)  [unwired: 9 in, 1 out]
            n540 = call "从动态数据转换47"("Dynamic Data Type"=w921) -> ("Array"=→"1609 7":dbl[])  [unwired: 3 in]
          }
        }
        n541 = case shown="1" w727 {
          tunnel: w747 -> [_ w833 w838 w841 w844 w845 w850]
          frame -1, Default {
          }
          frame 0 {
            n542 = call "信号收集器67"("Signals"=w833) -> ("Collected Signals"=w834:dynamicdata)  [unwired: 9 in, 1 out]
            n543 = call "从动态数据转换73"("Dynamic Data Type"=w834) -> ("Array"=→"1050 9":dbl[])  [unwired: 3 in]
          }
          frame 1 {
            n544 = call "信号收集器68"("Signals"=w838) -> ("Collected Signals"=w836:dynamicdata)  [unwired: 9 in, 1 out]
            n545 = call "从动态数据转换74"("Dynamic Data Type"=w836) -> ("Array"=→"1213 9":dbl[])  [unwired: 3 in]
          }
          frame 2 {
            n546 = call "信号收集器69"("Signals"=w841) -> ("Collected Signals"=w840:dynamicdata)  [unwired: 9 in, 1 out]
            n547 = call "从动态数据转换75"("Dynamic Data Type"=w840) -> ("Array"=→"1314 9":dbl[])  [unwired: 3 in]
          }
          frame 3 {
            n548 = call "信号收集器70"("Signals"=w844) -> ("Collected Signals"=w843:dynamicdata)  [unwired: 9 in, 1 out]
            n549 = call "从动态数据转换76"("Dynamic Data Type"=w843) -> ("Array"=→"1409 9":dbl[])  [unwired: 3 in]
          }
          frame 4 {
            n550 = call "信号收集器71"("Signals"=w845) -> ("Collected Signals"=w847:dynamicdata)  [unwired: 9 in, 1 out]
            n551 = call "从动态数据转换71"("Dynamic Data Type"=w847) -> ("Array"=→"1550 45":dbl[])  [unwired: 3 in]
          }
          frame 5 {
            n552 = call "信号收集器72"("Signals"=w850) -> ("Collected Signals"=w848:dynamicdata)  [unwired: 9 in, 1 out]
            n553 = call "从动态数据转换72"("Dynamic Data Type"=w848) -> ("Array"=→"1609 9":dbl[])  [unwired: 3 in]
          }
        }
        n554 = case shown="0" w727 {
          tunnel: w771 -> [_ w923 w928 w931 w934 w935 w940]
          frame -1, Default {
          }
          frame 0 {
            n555 = call "信号收集器37"("Signals"=w923) -> ("Collected Signals"=w924:dynamicdata)  [unwired: 9 in, 1 out]
            n556 = call "从动态数据转换41"("Dynamic Data Type"=w924) -> ("Array"=→"1050 8":dbl[])  [unwired: 3 in]
          }
          frame 1 {
            n557 = call "信号收集器38"("Signals"=w928) -> ("Collected Signals"=w926:dynamicdata)  [unwired: 9 in, 1 out]
            n558 = call "从动态数据转换42"("Dynamic Data Type"=w926) -> ("Array"=→"1213 8":dbl[])  [unwired: 3 in]
          }
          frame 2 {
            n559 = call "信号收集器39"("Signals"=w931) -> ("Collected Signals"=w929:dynamicdata)  [unwired: 9 in, 1 out]
            n560 = call "从动态数据转换43"("Dynamic Data Type"=w929) -> ("Array"=→"1314 8":dbl[])  [unwired: 3 in]
          }
          frame 3 {
            n561 = call "信号收集器40"("Signals"=w934) -> ("Collected Signals"=w933:dynamicdata)  [unwired: 9 in, 1 out]
            n562 = call "从动态数据转换44"("Dynamic Data Type"=w933) -> ("Array"=→"1409 8":dbl[])  [unwired: 3 in]
          }
          frame 4 {
            n563 = call "信号收集器41"("Signals"=w935) -> ("Collected Signals"=w937:dynamicdata)  [unwired: 9 in, 1 out]
            n564 = call "从动态数据转换45"("Dynamic Data Type"=w937) -> ("Array"=→"1550 8":dbl[])  [unwired: 3 in]
          }
          frame 5 {
            n565 = call "信号收集器42"("Signals"=w940) -> ("Collected Signals"=w938:dynamicdata)  [unwired: 9 in, 1 out]
            n566 = call "从动态数据转换46"("Dynamic Data Type"=w938) -> ("Array"=→"1609 8":dbl[])  [unwired: 3 in]
          }
        }
        n567 = case shown="3" w727 {
          tunnel: w764 -> [_ w869 w874 w877 w880 w881 w884]
          frame -1, Default {
          }
          frame 0 {
            n568 = call "信号收集器55"("Signals"=w869) -> ("Collected Signals"=w871:dynamicdata)  [unwired: 9 in, 1 out]
            n569 = call "从动态数据转换61"("Dynamic Data Type"=w871) -> ("Array"=→"1050 11":dbl[])  [unwired: 3 in]
          }
          frame 1 {
            n570 = call "信号收集器56"("Signals"=w874) -> ("Collected Signals"=w873:dynamicdata)  [unwired: 9 in, 1 out]
            n571 = call "从动态数据转换62"("Dynamic Data Type"=w873) -> ("Array"=→"1213 11":dbl[])  [unwired: 3 in]
          }
          frame 2 {
            n572 = call "信号收集器57"("Signals"=w877) -> ("Collected Signals"=w876:dynamicdata)  [unwired: 9 in, 1 out]
            n573 = call "从动态数据转换63"("Dynamic Data Type"=w876) -> ("Array"=→"1314 11":dbl[])  [unwired: 3 in]
          }
          frame 3 {
            n574 = call "信号收集器58"("Signals"=w880) -> ("Collected Signals"=w879:dynamicdata)  [unwired: 9 in, 1 out]
            n575 = call "从动态数据转换64"("Dynamic Data Type"=w879) -> ("Array"=→"1409 11":dbl[])  [unwired: 3 in]
          }
          frame 4 {
            n576 = call "信号收集器59"("Signals"=w881) -> ("Collected Signals"=w883:dynamicdata)  [unwired: 9 in, 1 out]
            n577 = call "从动态数据转换59"("Dynamic Data Type"=w883) -> ("Array"=→"1550 11":dbl[])  [unwired: 3 in]
          }
          frame 5 {
            n578 = call "信号收集器60"("Signals"=w884) -> ("Collected Signals"=w886:dynamicdata)  [unwired: 9 in, 1 out]
            n579 = call "从动态数据转换60"("Dynamic Data Type"=w886) -> ("Array"=→"1609 11":dbl[])  [unwired: 3 in]
          }
        }
        n580 = case shown="1" w727 {
          tunnel: w762 -> [_ w889 w892 w895 w898 w901 w904]
          frame -1, Default {
          }
          frame 0 {
            n581 = call "信号收集器49"("Signals"=w889) -> ("Collected Signals"=w888:dynamicdata)  [unwired: 9 in, 1 out]
            n582 = call "从动态数据转换55"("Dynamic Data Type"=w888) -> ("Array"=→"1050 6":dbl[])  [unwired: 3 in]
          }
          frame 1 {
            n583 = call "信号收集器50"("Signals"=w892) -> ("Collected Signals"=w891:dynamicdata)  [unwired: 9 in, 1 out]
            n584 = call "从动态数据转换56"("Dynamic Data Type"=w891) -> ("Array"=→"1213 6":dbl[])  [unwired: 3 in]
          }
          frame 2 {
            n585 = call "信号收集器51"("Signals"=w895) -> ("Collected Signals"=w894:dynamicdata)  [unwired: 9 in, 1 out]
            n586 = call "从动态数据转换57"("Dynamic Data Type"=w894) -> ("Array"=→"1314 6":dbl[])  [unwired: 3 in]
          }
          frame 3 {
            n587 = call "信号收集器52"("Signals"=w898) -> ("Collected Signals"=w897:dynamicdata)  [unwired: 9 in, 1 out]
            n588 = call "从动态数据转换58"("Dynamic Data Type"=w897) -> ("Array"=→"1409 6":dbl[])  [unwired: 3 in]
          }
          frame 4 {
            n589 = call "信号收集器53"("Signals"=w901) -> ("Collected Signals"=w899:dynamicdata)  [unwired: 9 in, 1 out]
            n590 = call "从动态数据转换53"("Dynamic Data Type"=w899) -> ("Array"=→"1550 6":dbl[])  [unwired: 3 in]
          }
          frame 5 {
            n591 = call "信号收集器54"("Signals"=w904) -> ("Collected Signals"=w903:dynamicdata)  [unwired: 9 in, 1 out]
            n592 = call "从动态数据转换54"("Dynamic Data Type"=w903) -> ("Array"=→"1609 6":dbl[])  [unwired: 3 in]
          }
        }
        n593 = case shown="1" w727 {
          tunnel: w758 -> [_ w815 w820 w821 w826 w827 w832]
          frame -1, Default {
          }
          frame 0 {
            n594 = call "信号收集器73"("Signals"=w815) -> ("Collected Signals"=w817:dynamicdata)  [unwired: 9 in, 1 out]
            n595 = call "从动态数据转换77"("Dynamic Data Type"=w817) -> ("Array"=→"1050 14":dbl[])  [unwired: 3 in]
          }
          frame 1 {
            n596 = call "信号收集器74"("Signals"=w820) -> ("Collected Signals"=w818:dynamicdata)  [unwired: 9 in, 1 out]
            n597 = call "从动态数据转换78"("Dynamic Data Type"=w818) -> ("Array"=→"1213 14":dbl[])  [unwired: 3 in]
          }
          frame 2 {
            n598 = call "信号收集器75"("Signals"=w821) -> ("Collected Signals"=w822:dynamicdata)  [unwired: 9 in, 1 out]
            n599 = call "从动态数据转换79"("Dynamic Data Type"=w822) -> ("Array"=→"1314 14":dbl[])  [unwired: 3 in]
          }
          frame 3 {
            n600 = call "信号收集器76"("Signals"=w826) -> ("Collected Signals"=w825:dynamicdata)  [unwired: 9 in, 1 out]
            n601 = call "从动态数据转换80"("Dynamic Data Type"=w825) -> ("Array"=→"1409 14":dbl[])  [unwired: 3 in]
          }
          frame 4 {
            n602 = call "信号收集器77"("Signals"=w827) -> ("Collected Signals"=w828:dynamicdata)  [unwired: 9 in, 1 out]
            n603 = call "从动态数据转换81"("Dynamic Data Type"=w828) -> ("Array"=→"1550 24":dbl[])  [unwired: 3 in]
          }
          frame 5 {
            n604 = call "信号收集器78"("Signals"=w832) -> ("Collected Signals"=w830:dynamicdata)  [unwired: 9 in, 1 out]
            n605 = call "从动态数据转换82"("Dynamic Data Type"=w830) -> ("Array"=→"1609 14":dbl[])  [unwired: 3 in]
          }
        }
        n606 = case shown="5" w727 {
          tunnel: w756 -> [_ w779 w784 w787 w790 w791 w796]
          frame -1, Default {
          }
          frame 0 {
            n607 = call "信号收集器85"("Signals"=w779) -> ("Collected Signals"=w781:dynamicdata)  [unwired: 9 in, 1 out]
            n608 = call "从动态数据转换92"("Dynamic Data Type"=w781) -> ("Array"=→"1050 12":dbl[])  [unwired: 3 in]
          }
          frame 1 {
            n609 = call "信号收集器86"("Signals"=w784) -> ("Collected Signals"=w783:dynamicdata)  [unwired: 9 in, 1 out]
            n610 = call "从动态数据转换93"("Dynamic Data Type"=w783) -> ("Array"=→"1213 12":dbl[])  [unwired: 3 in]
          }
          frame 2 {
            n611 = call "信号收集器87"("Signals"=w787) -> ("Collected Signals"=w786:dynamicdata)  [unwired: 9 in, 1 out]
            n612 = call "从动态数据转换94"("Dynamic Data Type"=w786) -> ("Array"=→"1314 12":dbl[])  [unwired: 3 in]
          }
          frame 3 {
            n613 = call "信号收集器88"("Signals"=w790) -> ("Collected Signals"=w789:dynamicdata)  [unwired: 9 in, 1 out]
            n614 = call "从动态数据转换87"("Dynamic Data Type"=w789) -> ("Array"=→"1409 12":dbl[])  [unwired: 3 in]
          }
          frame 4 {
            n615 = call "信号收集器89"("Signals"=w791) -> ("Collected Signals"=w792:dynamicdata)  [unwired: 9 in, 1 out]
            n616 = call "从动态数据转换90"("Dynamic Data Type"=w792) -> ("Array"=→"1550 12":dbl[])  [unwired: 3 in]
          }
          frame 5 {
            n617 = call "信号收集器90"("Signals"=w796) -> ("Collected Signals"=w795:dynamicdata)  [unwired: 9 in, 1 out]
            n618 = call "从动态数据转换91"("Dynamic Data Type"=w795) -> ("Array"=→"1609 12":dbl[])  [unwired: 3 in]
          }
        }
        n619 = call <vilib>:"Add State(s) to Queue__JKI_lib_State_Machine.vi"("State(s) in (\"\")"=w778) -> ("States Out"=w777:string)  [unwired: 14 in]
      }
      frame "UI: Update Graph_Diff_7R" {
        (unwired) 20 ("索引")
        (unwired) 19 ("索引")
        (unwired) 18 ("索引")
        (unwired) 17 ("索引")
        (unwired) 16 ("索引")
        (unwired) 15 ("索引")
        (unwired) 14 ("索引")
        (unwired) 13 ("索引")
        (unwired) 12 ("索引")
        (unwired) 11 ("索引")
        (unwired) 10 ("索引")
        # "短期-差分7环"
        # "5-7"
        # "6-7"
        # "5-6"
        # "4-6"
        # "4-7"
        # "3-6"
        # "3-7"
        # "2-6"
        # "2-7"
        # "1-6"
        # "1-7"
        # "#CSM \"Category Seperator\"\nDo not put any code in this frame."
        n620 = Unbundle By Name(w1061) -> ("Time and Data.当前运行信息.当前索引子集"=w1062:i8[], "Time and Data.Data"=w1070:dbl[], "Sample Settings.校准.温度校准值"=w1060:dbl[])
        n621 = Index Array(array=w1062) -> (element=w1059:i8)  [unwired: 1 in]
        n622 = Index Array(array=w1070) -> (element #1=w1067:dbl, element #2=w1066:dbl, element #3=w1065:dbl, element #4=w1064:dbl, element #5=w1063:dbl, element #6=w1069:dbl, element #7=w1068:dbl)  [unwired: 7 in]
        n623 = xnode "公式 16"("X1"=w1067, "X2"=w1069) -> ("结果"=w1101:dbl)  [unwired: 1 in, 1 out]
        n624 = xnode "公式 17"("X1"=w1067, "X2"=w1068) -> ("结果"=w1103:dbl)  [unwired: 1 in, 1 out]
        n625 = xnode "公式 26"("X1"=w1066, "X2"=w1069) -> ("结果"=w1095:dbl)  [unwired: 1 in, 1 out]
        n626 = xnode "公式 27"("X1"=w1066, "X2"=w1068) -> ("结果"=w1097:dbl)  [unwired: 1 in, 1 out]
        n627 = xnode "公式 36"("X1"=w1065, "X2"=w1069) -> ("结果"=w1089:dbl)  [unwired: 1 in, 1 out]
        n628 = xnode "公式 37"("X1"=w1065, "X2"=w1068) -> ("结果"=w1091:dbl)  [unwired: 1 in, 1 out]
        n629 = xnode "公式 46"("X1"=w1064, "X2"=w1069) -> ("结果"=w1083:dbl)  [unwired: 1 in, 1 out]
        n630 = xnode "公式 47"("X1"=w1064, "X2"=w1068) -> ("结果"=w1085:dbl)  [unwired: 1 in, 1 out]
        n631 = xnode "公式 56"("X1"=w1063, "X2"=w1069) -> ("结果"=w1079:dbl)  [unwired: 1 in, 1 out]
        n632 = xnode "公式 57"("X1"=w1063, "X2"=w1068) -> ("结果"=w1074:dbl)  [unwired: 1 in, 1 out]
        n633 = xnode "公式 67"("X1"=w1069, "X2"=w1068) -> ("结果"=w1076:dbl)  [unwired: 1 in, 1 out]
        n634 = Index Array(array=w1060) -> (element=w1102:dbl)  [unwired: 1 in]
        n635 = Index Array(array=w1060) -> (element=w1096:dbl)  [unwired: 1 in]
        n636 = Index Array(array=w1060) -> (element=w1090:dbl)  [unwired: 1 in]
        n637 = Index Array(array=w1060) -> (element=w1084:dbl)  [unwired: 1 in]
        n638 = Index Array(array=w1060) -> (element=w1078:dbl)  [unwired: 1 in]
        n639 = Index Array(array=w1060) -> (element=w1075:dbl)  [unwired: 1 in]
        n640 = Index Array(array=w1060) -> (element=w1100:dbl)  [unwired: 1 in]
        n641 = Index Array(array=w1060) -> (element=w1094:dbl)  [unwired: 1 in]
        n642 = Index Array(array=w1060) -> (element=w1088:dbl)  [unwired: 1 in]
        n643 = Index Array(array=w1060) -> (element=w1082:dbl)  [unwired: 1 in]
        n644 = Index Array(array=w1060) -> (element=w1073:dbl)  [unwired: 1 in]
        n645 = Subtract(x=w1103, y=w1102) -> (x-y=w1099:dbl)
        n646 = Subtract(x=w1097, y=w1096) -> (x-y=w1093:dbl)
        n647 = Subtract(x=w1091, y=w1090) -> (x-y=w1087:dbl)
        n648 = Subtract(x=w1085, y=w1084) -> (x-y=w1081:dbl)
        n649 = Subtract(x=w1079, y=w1078) -> (x-y=w1077:dbl)
        n650 = Subtract(x=w1076, y=w1075) -> (x-y=w1072:dbl)
        n651 = Subtract(x=w1101, y=w1100) -> (x-y=w1098:dbl)
        n652 = Subtract(x=w1095, y=w1094) -> (x-y=w1092:dbl)
        n653 = Subtract(x=w1089, y=w1088) -> (x-y=w1086:dbl)
        n654 = Subtract(x=w1083, y=w1082) -> (x-y=w1080:dbl)
        n655 = Subtract(x=w1074, y=w1073) -> (x-y=w1071:dbl)
        n656 = case shown="3" w1059 {
          tunnel: w1099 -> [_ w1379 w1383 w1386 w1389 w1391 w1395]
          frame -1, Default {
          }
          frame 0 {
            n657 = call "信号收集器109"("Signals"=w1379) -> ("Collected Signals"=w1380:dynamicdata)  [unwired: 9 in, 1 out]
            n658 = call "从动态数据转换109"("Dynamic Data Type"=w1380) -> ("Array"=→"1050 19":dbl[])  [unwired: 3 in]
          }
          frame 1 {
            n659 = call "信号收集器110"("Signals"=w1383) -> ("Collected Signals"=w1382:dynamicdata)  [unwired: 9 in, 1 out]
            n660 = call "从动态数据转换110"("Dynamic Data Type"=w1382) -> ("Array"=→"1213 19":dbl[])  [unwired: 3 in]
          }
          frame 2 {
            n661 = call "信号收集器111"("Signals"=w1386) -> ("Collected Signals"=w1385:dynamicdata)  [unwired: 9 in, 1 out]
            n662 = call "从动态数据转换111"("Dynamic Data Type"=w1385) -> ("Array"=→"1314 19":dbl[])  [unwired: 3 in]
          }
          frame 3 {
            n663 = call "信号收集器112"("Signals"=w1389) -> ("Collected Signals"=w1388:dynamicdata)  [unwired: 9 in, 1 out]
            n664 = call "从动态数据转换112"("Dynamic Data Type"=w1388) -> ("Array"=→"1409 19":dbl[])  [unwired: 3 in]
          }
          frame 4 {
            n665 = call "信号收集器113"("Signals"=w1391) -> ("Collected Signals"=w1392:dynamicdata)  [unwired: 9 in, 1 out]
            n666 = call "从动态数据转换113"("Dynamic Data Type"=w1392) -> ("Array"=→"1550 17":dbl[])  [unwired: 3 in]
          }
          frame 5 {
            n667 = call "信号收集器114"("Signals"=w1395) -> ("Collected Signals"=w1394:dynamicdata)  [unwired: 9 in, 1 out]
            n668 = call "从动态数据转换114"("Dynamic Data Type"=w1394) -> ("Array"=→"1609 19":dbl[])  [unwired: 3 in]
          }
        }
        n669 = case shown="0" w1059 {
          tunnel: w1093 -> [_ w1323 w1327 w1330 w1333 w1335 w1339]
          frame -1, Default {
          }
          frame 0 {
            n670 = call "信号收集器121"("Signals"=w1323) -> ("Collected Signals"=w1324:dynamicdata)  [unwired: 9 in, 1 out]
            n671 = call "从动态数据转换121"("Dynamic Data Type"=w1324) -> ("Array"=→"1050 21":dbl[])  [unwired: 3 in]
          }
          frame 1 {
            n672 = call "信号收集器122"("Signals"=w1327) -> ("Collected Signals"=w1326:dynamicdata)  [unwired: 9 in, 1 out]
            n673 = call "从动态数据转换122"("Dynamic Data Type"=w1326) -> ("Array"=→"1213 21":dbl[])  [unwired: 3 in]
          }
          frame 2 {
            n674 = call "信号收集器123"("Signals"=w1330) -> ("Collected Signals"=w1329:dynamicdata)  [unwired: 9 in, 1 out]
            n675 = call "从动态数据转换123"("Dynamic Data Type"=w1329) -> ("Array"=→"1314 21":dbl[])  [unwired: 3 in]
          }
          frame 3 {
            n676 = call "信号收集器124"("Signals"=w1333) -> ("Collected Signals"=w1332:dynamicdata)  [unwired: 9 in, 1 out]
            n677 = call "从动态数据转换124"("Dynamic Data Type"=w1332) -> ("Array"=→"1409 21":dbl[])  [unwired: 3 in]
          }
          frame 4 {
            n678 = call "信号收集器125"("Signals"=w1335) -> ("Collected Signals"=w1336:dynamicdata)  [unwired: 9 in, 1 out]
            n679 = call "从动态数据转换125"("Dynamic Data Type"=w1336) -> ("Array"=→"1550 19":dbl[])  [unwired: 3 in]
          }
          frame 5 {
            n680 = call "信号收集器126"("Signals"=w1339) -> ("Collected Signals"=w1338:dynamicdata)  [unwired: 9 in, 1 out]
            n681 = call "从动态数据转换126"("Dynamic Data Type"=w1338) -> ("Array"=→"1609 21":dbl[])  [unwired: 3 in]
          }
        }
        n682 = case shown="0" w1059 {
          tunnel: w1087 -> [_ w1267 w1271 w1274 w1277 w1279 w1283]
          frame -1, Default {
          }
          frame 0 {
            n683 = call "信号收集器133"("Signals"=w1267) -> ("Collected Signals"=w1268:dynamicdata)  [unwired: 9 in, 1 out]
            n684 = call "从动态数据转换133"("Dynamic Data Type"=w1268) -> ("Array"=→"1050 23":dbl[])  [unwired: 3 in]
          }
          frame 1 {
            n685 = call "信号收集器134"("Signals"=w1271) -> ("Collected Signals"=w1270:dynamicdata)  [unwired: 9 in, 1 out]
            n686 = call "从动态数据转换134"("Dynamic Data Type"=w1270) -> ("Array"=→"1213 23":dbl[])  [unwired: 3 in]
          }
          frame 2 {
            n687 = call "信号收集器135"("Signals"=w1274) -> ("Collected Signals"=w1273:dynamicdata)  [unwired: 9 in, 1 out]
            n688 = call "从动态数据转换135"("Dynamic Data Type"=w1273) -> ("Array"=→"1314 23":dbl[])  [unwired: 3 in]
          }
          frame 3 {
            n689 = call "信号收集器136"("Signals"=w1277) -> ("Collected Signals"=w1276:dynamicdata)  [unwired: 9 in, 1 out]
            n690 = call "从动态数据转换136"("Dynamic Data Type"=w1276) -> ("Array"=→"1409 23":dbl[])  [unwired: 3 in]
          }
          frame 4 {
            n691 = call "信号收集器137"("Signals"=w1279) -> ("Collected Signals"=w1280:dynamicdata)  [unwired: 9 in, 1 out]
            n692 = call "从动态数据转换137"("Dynamic Data Type"=w1280) -> ("Array"=→"1550 21":dbl[])  [unwired: 3 in]
          }
          frame 5 {
            n693 = call "信号收集器138"("Signals"=w1283) -> ("Collected Signals"=w1282:dynamicdata)  [unwired: 9 in, 1 out]
            n694 = call "从动态数据转换138"("Dynamic Data Type"=w1282) -> ("Array"=→"1609 23":dbl[])  [unwired: 3 in]
          }
        }
        n695 = case shown="4" w1059 {
          tunnel: w1081 -> [_ w1211 w1215 w1218 w1221 w1223 w1227]
          frame -1, Default {
          }
          frame 0 {
            n696 = call "信号收集器145"("Signals"=w1211) -> ("Collected Signals"=w1212:dynamicdata)  [unwired: 9 in, 1 out]
            n697 = call "从动态数据转换145"("Dynamic Data Type"=w1212) -> ("Array"=→"1050 25":dbl[])  [unwired: 3 in]
          }
          frame 1 {
            n698 = call "信号收集器146"("Signals"=w1215) -> ("Collected Signals"=w1214:dynamicdata)  [unwired: 9 in, 1 out]
            n699 = call "从动态数据转换146"("Dynamic Data Type"=w1214) -> ("Array"=→"1213 25":dbl[])  [unwired: 3 in]
          }
          frame 2 {
            n700 = call "信号收集器147"("Signals"=w1218) -> ("Collected Signals"=w1217:dynamicdata)  [unwired: 9 in, 1 out]
            n701 = call "从动态数据转换147"("Dynamic Data Type"=w1217) -> ("Array"=→"1314 25":dbl[])  [unwired: 3 in]
          }
          frame 3 {
            n702 = call "信号收集器148"("Signals"=w1221) -> ("Collected Signals"=w1220:dynamicdata)  [unwired: 9 in, 1 out]
            n703 = call "从动态数据转换148"("Dynamic Data Type"=w1220) -> ("Array"=→"1409 25":dbl[])  [unwired: 3 in]
          }
          frame 4 {
            n704 = call "信号收集器149"("Signals"=w1223) -> ("Collected Signals"=w1224:dynamicdata)  [unwired: 9 in, 1 out]
            n705 = call "从动态数据转换149"("Dynamic Data Type"=w1224) -> ("Array"=→"1550 23":dbl[])  [unwired: 3 in]
          }
          frame 5 {
            n706 = call "信号收集器150"("Signals"=w1227) -> ("Collected Signals"=w1226:dynamicdata)  [unwired: 9 in, 1 out]
            n707 = call "从动态数据转换150"("Dynamic Data Type"=w1226) -> ("Array"=→"1609 25":dbl[])  [unwired: 3 in]
          }
        }
        n708 = case shown="0" w1059 {
          tunnel: w1077 -> [_ w1173 w1177 w1180 w1183 w1185 w1189]
          frame -1, Default {
          }
          frame 0 {
            n709 = call "信号收集器151"("Signals"=w1173) -> ("Collected Signals"=w1174:dynamicdata)  [unwired: 9 in, 1 out]
            n710 = call "从动态数据转换151"("Dynamic Data Type"=w1174) -> ("Array"=→"1050 26":dbl[])  [unwired: 3 in]
          }
          frame 1 {
            n711 = call "信号收集器152"("Signals"=w1177) -> ("Collected Signals"=w1176:dynamicdata)  [unwired: 9 in, 1 out]
            n712 = call "从动态数据转换152"("Dynamic Data Type"=w1176) -> ("Array"=→"1213 26":dbl[])  [unwired: 3 in]
          }
          frame 2 {
            n713 = call "信号收集器153"("Signals"=w1180) -> ("Collected Signals"=w1179:dynamicdata)  [unwired: 9 in, 1 out]
            n714 = call "从动态数据转换153"("Dynamic Data Type"=w1179) -> ("Array"=→"1314 26":dbl[])  [unwired: 3 in]
          }
          frame 3 {
            n715 = call "信号收集器154"("Signals"=w1183) -> ("Collected Signals"=w1182:dynamicdata)  [unwired: 9 in, 1 out]
            n716 = call "从动态数据转换154"("Dynamic Data Type"=w1182) -> ("Array"=→"1409 26":dbl[])  [unwired: 3 in]
          }
          frame 4 {
            n717 = call "信号收集器155"("Signals"=w1185) -> ("Collected Signals"=w1186:dynamicdata)  [unwired: 9 in, 1 out]
            n718 = call "从动态数据转换155"("Dynamic Data Type"=w1186) -> ("Array"=→"1550 25":dbl[])  [unwired: 3 in]
          }
          frame 5 {
            n719 = call "信号收集器156"("Signals"=w1189) -> ("Collected Signals"=w1188:dynamicdata)  [unwired: 9 in, 1 out]
            n720 = call "从动态数据转换156"("Dynamic Data Type"=w1188) -> ("Array"=→"1609 26":dbl[])  [unwired: 3 in]
          }
        }
        n721 = case shown="5" w1059 {
          tunnel: w1098 -> [_ w1397 w1401 w1404 w1407 w1409 w1413]
          frame -1, Default {
          }
          frame 0 {
            n722 = call "信号收集器103"("Signals"=w1397) -> ("Collected Signals"=w1398:dynamicdata)  [unwired: 9 in, 1 out]
            n723 = call "从动态数据转换103"("Dynamic Data Type"=w1398) -> ("Array"=→"1050 18":dbl[])  [unwired: 3 in]
          }
          frame 1 {
            n724 = call "信号收集器104"("Signals"=w1401) -> ("Collected Signals"=w1400:dynamicdata)  [unwired: 9 in, 1 out]
            n725 = call "从动态数据转换104"("Dynamic Data Type"=w1400) -> ("Array"=→"1213 18":dbl[])  [unwired: 3 in]
          }
          frame 2 {
            n726 = call "信号收集器105"("Signals"=w1404) -> ("Collected Signals"=w1403:dynamicdata)  [unwired: 9 in, 1 out]
            n727 = call "从动态数据转换105"("Dynamic Data Type"=w1403) -> ("Array"=→"1314 18":dbl[])  [unwired: 3 in]
          }
          frame 3 {
            n728 = call "信号收集器106"("Signals"=w1407) -> ("Collected Signals"=w1406:dynamicdata)  [unwired: 9 in, 1 out]
            n729 = call "从动态数据转换106"("Dynamic Data Type"=w1406) -> ("Array"=→"1409 18":dbl[])  [unwired: 3 in]
          }
          frame 4 {
            n730 = call "信号收集器107"("Signals"=w1409) -> ("Collected Signals"=w1410:dynamicdata)  [unwired: 9 in, 1 out]
            n731 = call "从动态数据转换107"("Dynamic Data Type"=w1410) -> ("Array"=→"1550 16":dbl[])  [unwired: 3 in]
          }
          frame 5 {
            n732 = call "信号收集器108"("Signals"=w1413) -> ("Collected Signals"=w1412:dynamicdata)  [unwired: 9 in, 1 out]
            n733 = call "从动态数据转换108"("Dynamic Data Type"=w1412) -> ("Array"=→"1609 18":dbl[])  [unwired: 3 in]
          }
        }
        n734 = case shown="3" w1059 {
          tunnel: w1092 -> [_ w1341 w1345 w1348 w1351 w1353 w1357]
          frame -1, Default {
          }
          frame 0 {
            n735 = call "信号收集器115"("Signals"=w1341) -> ("Collected Signals"=w1342:dynamicdata)  [unwired: 9 in, 1 out]
            n736 = call "从动态数据转换115"("Dynamic Data Type"=w1342) -> ("Array"=→"1050 20":dbl[])  [unwired: 3 in]
          }
          frame 1 {
            n737 = call "信号收集器116"("Signals"=w1345) -> ("Collected Signals"=w1344:dynamicdata)  [unwired: 9 in, 1 out]
            n738 = call "从动态数据转换116"("Dynamic Data Type"=w1344) -> ("Array"=→"1213 20":dbl[])  [unwired: 3 in]
          }
          frame 2 {
            n739 = call "信号收集器117"("Signals"=w1348) -> ("Collected Signals"=w1347:dynamicdata)  [unwired: 9 in, 1 out]
            n740 = call "从动态数据转换117"("Dynamic Data Type"=w1347) -> ("Array"=→"1314 20":dbl[])  [unwired: 3 in]
          }
          frame 3 {
            n741 = call "信号收集器118"("Signals"=w1351) -> ("Collected Signals"=w1350:dynamicdata)  [unwired: 9 in, 1 out]
            n742 = call "从动态数据转换118"("Dynamic Data Type"=w1350) -> ("Array"=→"1409 20":dbl[])  [unwired: 3 in]
          }
          frame 4 {
            n743 = call "信号收集器119"("Signals"=w1353) -> ("Collected Signals"=w1354:dynamicdata)  [unwired: 9 in, 1 out]
            n744 = call "从动态数据转换119"("Dynamic Data Type"=w1354) -> ("Array"=→"1550 18":dbl[])  [unwired: 3 in]
          }
          frame 5 {
            n745 = call "信号收集器120"("Signals"=w1357) -> ("Collected Signals"=w1356:dynamicdata)  [unwired: 9 in, 1 out]
            n746 = call "从动态数据转换120"("Dynamic Data Type"=w1356) -> ("Array"=→"1609 20":dbl[])  [unwired: 3 in]
          }
        }
        n747 = case shown="1" w1059 {
          tunnel: w1072 -> [_ w1127 w1131 w1134 w1137 w1139 w1143]
          frame -1, Default {
          }
          frame 0 {
            n748 = call "信号收集器163"("Signals"=w1127) -> ("Collected Signals"=w1128:dynamicdata)  [unwired: 9 in, 1 out]
            n749 = call "从动态数据转换163"("Dynamic Data Type"=w1128) -> ("Array"=→"1050 17":dbl[])  [unwired: 3 in]
          }
          frame 1 {
            n750 = call "信号收集器164"("Signals"=w1131) -> ("Collected Signals"=w1130:dynamicdata)  [unwired: 9 in, 1 out]
            n751 = call "从动态数据转换164"("Dynamic Data Type"=w1130) -> ("Array"=→"1213 17":dbl[])  [unwired: 3 in]
          }
          frame 2 {
            n752 = call "信号收集器165"("Signals"=w1134) -> ("Collected Signals"=w1133:dynamicdata)  [unwired: 9 in, 1 out]
            n753 = call "从动态数据转换165"("Dynamic Data Type"=w1133) -> ("Array"=→"1314 17":dbl[])  [unwired: 3 in]
          }
          frame 3 {
            n754 = call "信号收集器166"("Signals"=w1137) -> ("Collected Signals"=w1136:dynamicdata)  [unwired: 9 in, 1 out]
            n755 = call "从动态数据转换166"("Dynamic Data Type"=w1136) -> ("Array"=→"1409 17":dbl[])  [unwired: 3 in]
          }
          frame 4 {
            n756 = call "信号收集器167"("Signals"=w1139) -> ("Collected Signals"=w1140:dynamicdata)  [unwired: 9 in, 1 out]
            n757 = call "从动态数据转换167"("Dynamic Data Type"=w1140) -> ("Array"=→"1550 15":dbl[])  [unwired: 3 in]
          }
          frame 5 {
            n758 = call "信号收集器168"("Signals"=w1143) -> ("Collected Signals"=w1142:dynamicdata)  [unwired: 9 in, 1 out]
            n759 = call "从动态数据转换168"("Dynamic Data Type"=w1142) -> ("Array"=→"1609 17":dbl[])  [unwired: 3 in]
          }
        }
        n760 = case shown="0" w1059 {
          tunnel: w1086 -> [_ w1285 w1289 w1292 w1295 w1297 w1301]
          frame -1, Default {
          }
          frame 0 {
            n761 = call "信号收集器127"("Signals"=w1285) -> ("Collected Signals"=w1286:dynamicdata)  [unwired: 9 in, 1 out]
            n762 = call "从动态数据转换127"("Dynamic Data Type"=w1286) -> ("Array"=→"1050 22":dbl[])  [unwired: 3 in]
          }
          frame 1 {
            n763 = call "信号收集器128"("Signals"=w1289) -> ("Collected Signals"=w1288:dynamicdata)  [unwired: 9 in, 1 out]
            n764 = call "从动态数据转换128"("Dynamic Data Type"=w1288) -> ("Array"=→"1213 22":dbl[])  [unwired: 3 in]
          }
          frame 2 {
            n765 = call "信号收集器129"("Signals"=w1292) -> ("Collected Signals"=w1291:dynamicdata)  [unwired: 9 in, 1 out]
            n766 = call "从动态数据转换129"("Dynamic Data Type"=w1291) -> ("Array"=→"1314 22":dbl[])  [unwired: 3 in]
          }
          frame 3 {
            n767 = call "信号收集器130"("Signals"=w1295) -> ("Collected Signals"=w1294:dynamicdata)  [unwired: 9 in, 1 out]
            n768 = call "从动态数据转换130"("Dynamic Data Type"=w1294) -> ("Array"=→"1409 22":dbl[])  [unwired: 3 in]
          }
          frame 4 {
            n769 = call "信号收集器131"("Signals"=w1297) -> ("Collected Signals"=w1298:dynamicdata)  [unwired: 9 in, 1 out]
            n770 = call "从动态数据转换131"("Dynamic Data Type"=w1298) -> ("Array"=→"1550 20":dbl[])  [unwired: 3 in]
          }
          frame 5 {
            n771 = call "信号收集器132"("Signals"=w1301) -> ("Collected Signals"=w1300:dynamicdata)  [unwired: 9 in, 1 out]
            n772 = call "从动态数据转换132"("Dynamic Data Type"=w1300) -> ("Array"=→"1609 22":dbl[])  [unwired: 3 in]
          }
        }
        n773 = case shown="4" w1059 {
          tunnel: w1080 -> [_ w1229 w1233 w1236 w1239 w1241 w1245]
          frame -1, Default {
          }
          frame 0 {
            n774 = call "信号收集器139"("Signals"=w1229) -> ("Collected Signals"=w1230:dynamicdata)  [unwired: 9 in, 1 out]
            n775 = call "从动态数据转换139"("Dynamic Data Type"=w1230) -> ("Array"=→"1050 24":dbl[])  [unwired: 3 in]
          }
          frame 1 {
            n776 = call "信号收集器140"("Signals"=w1233) -> ("Collected Signals"=w1232:dynamicdata)  [unwired: 9 in, 1 out]
            n777 = call "从动态数据转换140"("Dynamic Data Type"=w1232) -> ("Array"=→"1213 24":dbl[])  [unwired: 3 in]
          }
          frame 2 {
            n778 = call "信号收集器141"("Signals"=w1236) -> ("Collected Signals"=w1235:dynamicdata)  [unwired: 9 in, 1 out]
            n779 = call "从动态数据转换141"("Dynamic Data Type"=w1235) -> ("Array"=→"1314 24":dbl[])  [unwired: 3 in]
          }
          frame 3 {
            n780 = call "信号收集器142"("Signals"=w1239) -> ("Collected Signals"=w1238:dynamicdata)  [unwired: 9 in, 1 out]
            n781 = call "从动态数据转换142"("Dynamic Data Type"=w1238) -> ("Array"=→"1409 24":dbl[])  [unwired: 3 in]
          }
          frame 4 {
            n782 = call "信号收集器143"("Signals"=w1241) -> ("Collected Signals"=w1242:dynamicdata)  [unwired: 9 in, 1 out]
            n783 = call "从动态数据转换143"("Dynamic Data Type"=w1242) -> ("Array"=→"1550 22":dbl[])  [unwired: 3 in]
          }
          frame 5 {
            n784 = call "信号收集器144"("Signals"=w1245) -> ("Collected Signals"=w1244:dynamicdata)  [unwired: 9 in, 1 out]
            n785 = call "从动态数据转换144"("Dynamic Data Type"=w1244) -> ("Array"=→"1609 24":dbl[])  [unwired: 3 in]
          }
        }
        n786 = case shown="4" w1059 {
          tunnel: w1071 -> [_ w1145 w1149 w1152 w1155 w1157 w1161]
          frame -1, Default {
          }
          frame 0 {
            n787 = call "信号收集器157"("Signals"=w1145) -> ("Collected Signals"=w1146:dynamicdata)  [unwired: 9 in, 1 out]
            n788 = call "从动态数据转换157"("Dynamic Data Type"=w1146) -> ("Array"=→"1050 27":dbl[])  [unwired: 3 in]
          }
          frame 1 {
            n789 = call "信号收集器158"("Signals"=w1149) -> ("Collected Signals"=w1148:dynamicdata)  [unwired: 9 in, 1 out]
            n790 = call "从动态数据转换158"("Dynamic Data Type"=w1148) -> ("Array"=→"1213 27":dbl[])  [unwired: 3 in]
          }
          frame 2 {
            n791 = call "信号收集器159"("Signals"=w1152) -> ("Collected Signals"=w1151:dynamicdata)  [unwired: 9 in, 1 out]
            n792 = call "从动态数据转换159"("Dynamic Data Type"=w1151) -> ("Array"=→"1314 27":dbl[])  [unwired: 3 in]
          }
          frame 3 {
            n793 = call "信号收集器160"("Signals"=w1155) -> ("Collected Signals"=w1154:dynamicdata)  [unwired: 9 in, 1 out]
            n794 = call "从动态数据转换160"("Dynamic Data Type"=w1154) -> ("Array"=→"1409 27":dbl[])  [unwired: 3 in]
          }
          frame 4 {
            n795 = call "信号收集器161"("Signals"=w1157) -> ("Collected Signals"=w1158:dynamicdata)  [unwired: 9 in, 1 out]
            n796 = call "从动态数据转换161"("Dynamic Data Type"=w1158) -> ("Array"=→"1550 26":dbl[])  [unwired: 3 in]
          }
          frame 5 {
            n797 = call "信号收集器162"("Signals"=w1161) -> ("Collected Signals"=w1160:dynamicdata)  [unwired: 9 in, 1 out]
            n798 = call "从动态数据转换162"("Dynamic Data Type"=w1160) -> ("Array"=→"1609 27":dbl[])  [unwired: 3 in]
          }
        }
        n799 = call <vilib>:"Add State(s) to Queue__JKI_lib_State_Machine.vi"("State(s) in (\"\")"=w1105) -> ("States Out"=w1104:string)  [unwired: 14 in]
      }
      frame "UI: Update Graph_Single_LT" {
        # "长期-单环"
        n800 = Unbundle By Name(w1425) -> ("Time and Data.当前运行信息.当前索引子集"=w1424:i8[], "Indicators.图表相关.分段颜色"=w1416:enum32{"蓝色", "红色"}, "Time and Data.Data"=w1426:dbl[], "Indicators.图表相关.基准索引"=w1414:i32)
        n801 = Index Array(array=w1424) -> (element=w1415:i8)  [unwired: 1 in]
        n802 = Index Array(array=w1426) -> (element #1=w1423:dbl, element #2=w1422:dbl, element #3=w1421:dbl, element #4=w1420:dbl, element #5=w1419:dbl, element #6=w1418:dbl, element #7=w1417:dbl)  [unwired: 7 in]
        n803 = case shown="6" "单环Ca" {
          tunnel: w1423 -> [w1480 _ _ _ _ _ _]
          tunnel: w1422 -> [_ w1481 _ _ _ _ _]
          tunnel: w1421 -> [_ _ w1482 _ _ _ _]
          tunnel: w1420 -> [_ _ _ w1483 _ _ _]
          tunnel: [w1480 w1481 w1482 w1483 w1484 w1485 w1486] -> w1436
          tunnel: w1419 -> [_ _ _ _ w1484 _ _]
          tunnel: w1418 -> [_ _ _ _ _ w1485 _]
          tunnel: w1417 -> [_ _ _ _ _ _ w1486]
          frame 0, Default {
          }
          frame 1 {
          }
          frame 2 {
          }
          frame 3 {
          }
          frame 4 {
          }
          frame 5 {
          }
          frame 6 {
          }
        }
        n804 = case shown="0, 默认" "单环Aa" {
          tunnel: w1423 -> [w1522 _ _ _ _ _ _]
          tunnel: w1422 -> [_ w1523 _ _ _ _ _]
          tunnel: w1421 -> [_ _ w1524 _ _ _ _]
          tunnel: w1420 -> [_ _ _ w1525 _ _ _]
          tunnel: [w1522 w1523 w1524 w1525 w1526 w1527 w1528] -> w1445
          tunnel: w1419 -> [_ _ _ _ w1526 _ _]
          tunnel: w1418 -> [_ _ _ _ _ w1527 _]
          tunnel: w1417 -> [_ _ _ _ _ _ w1528]
          frame 0, Default {
          }
          frame 1 {
          }
          frame 2 {
          }
          frame 3 {
          }
          frame 4 {
          }
          frame 5 {
          }
          frame 6 {
          }
        }
        n805 = case shown="6" "单环Ba" {
          tunnel: w1423 -> [w1571 _ _ _ _ _ _]
          tunnel: w1422 -> [_ w1572 _ _ _ _ _]
          tunnel: w1421 -> [_ _ w1573 _ _ _ _]
          tunnel: w1420 -> [_ _ _ w1574 _ _ _]
          tunnel: [w1571 w1572 w1573 w1574 w1575 w1576 w1577] -> w1454
          tunnel: w1419 -> [_ _ _ _ w1575 _ _]
          tunnel: w1418 -> [_ _ _ _ _ w1576 _]
          tunnel: w1417 -> [_ _ _ _ _ _ w1577]
          frame 0, Default {
          }
          frame 1 {
          }
          frame 2 {
          }
          frame 3 {
          }
          frame 4 {
          }
          frame 5 {
          }
          frame 6 {
          }
        }
        n806 = case shown="6" "单环Cb" {
          tunnel: w1423 -> [w1473 _ _ _ _ _ _]
          tunnel: w1422 -> [_ w1474 _ _ _ _ _]
          tunnel: w1421 -> [_ _ w1475 _ _ _ _]
          tunnel: w1420 -> [_ _ _ w1476 _ _ _]
          tunnel: [w1473 w1474 w1475 w1476 w1477 w1478 w1479] -> w1437
          tunnel: w1419 -> [_ _ _ _ w1477 _ _]
          tunnel: w1418 -> [_ _ _ _ _ w1478 _]
          tunnel: w1417 -> [_ _ _ _ _ _ w1479]
          frame 0, Default {
          }
          frame 1 {
          }
          frame 2 {
          }
          frame 3 {
          }
          frame 4 {
          }
          frame 5 {
          }
          frame 6 {
          }
        }
        n807 = case shown="6" "单环Cc" {
          tunnel: w1423 -> [w1466 _ _ _ _ _ _]
          tunnel: w1422 -> [_ w1467 _ _ _ _ _]
          tunnel: w1421 -> [_ _ w1468 _ _ _ _]
          tunnel: w1420 -> [_ _ _ w1469 _ _ _]
          tunnel: [w1466 w1467 w1468 w1469 w1470 w1471 w1472] -> w1438
          tunnel: w1419 -> [_ _ _ _ w1470 _ _]
          tunnel: w1418 -> [_ _ _ _ _ w1471 _]
          tunnel: w1417 -> [_ _ _ _ _ _ w1472]
          frame 0, Default {
          }
          frame 1 {
          }
          frame 2 {
          }
          frame 3 {
          }
          frame 4 {
          }
          frame 5 {
          }
          frame 6 {
          }
        }
        n808 = case shown="5" "单环Ab" {
          tunnel: w1423 -> [w1529 _ _ _ _ _ _]
          tunnel: w1422 -> [_ w1530 _ _ _ _ _]
          tunnel: w1421 -> [_ _ w1531 _ _ _ _]
          tunnel: w1420 -> [_ _ _ w1532 _ _ _]
          tunnel: [w1529 w1530 w1531 w1532 w1533 w1534 w1535] -> w1446
          tunnel: w1419 -> [_ _ _ _ w1533 _ _]
          tunnel: w1418 -> [_ _ _ _ _ w1534 _]
          tunnel: w1417 -> [_ _ _ _ _ _ w1535]
          frame 0, Default {
          }
          frame 1 {
          }
          frame 2 {
          }
          frame 3 {
          }
          frame 4 {
          }
          frame 5 {
          }
          frame 6 {
          }
        }
        n809 = case shown="6" "单环Ac" {
          tunnel: w1423 -> [w1536 _ _ _ _ _ _]
          tunnel: w1422 -> [_ w1537 _ _ _ _ _]
          tunnel: w1421 -> [_ _ w1538 _ _ _ _]
          tunnel: w1420 -> [_ _ _ w1539 _ _ _]
          tunnel: [w1536 w1537 w1538 w1539 w1540 w1541 w1542] -> w1447
          tunnel: w1419 -> [_ _ _ _ w1540 _ _]
          tunnel: w1418 -> [_ _ _ _ _ w1541 _]
          tunnel: w1417 -> [_ _ _ _ _ _ w1542]
          tunnel: w1418 -> [_ _ _ _ _ _ _]
          tunnel: w1417 -> [_ _ _ _ _ _ _]
          frame 0, Default {
          }
          frame 1 {
          }
          frame 2 {
          }
          frame 3 {
          }
          frame 4 {
          }
          frame 5 {
          }
          frame 6 {
          }
        }
        n810 = case shown="6" "单环Bb" {
          tunnel: w1423 -> [w1564 _ _ _ _ _ _]
          tunnel: w1422 -> [_ w1565 _ _ _ _ _]
          tunnel: w1421 -> [_ _ w1566 _ _ _ _]
          tunnel: w1420 -> [_ _ _ w1567 _ _ _]
          tunnel: [w1564 w1565 w1566 w1567 w1568 w1569 w1570] -> w1453
          tunnel: w1419 -> [_ _ _ _ w1568 _ _]
          tunnel: w1418 -> [_ _ _ _ _ w1569 _]
          tunnel: w1417 -> [_ _ _ _ _ _ w1570]
          frame 0, Default {
          }
          frame 1 {
          }
          frame 2 {
          }
          frame 3 {
          }
          frame 4 {
          }
          frame 5 {
          }
          frame 6 {
          }
        }
        n811 = case shown="6" "单环Bc" {
          tunnel: w1423 -> [w1557 _ _ _ _ _ _]
          tunnel: w1422 -> [_ w1558 _ _ _ _ _]
          tunnel: w1421 -> [_ _ w1559 _ _ _ _]
          tunnel: w1420 -> [_ _ _ w1560 _ _ _]
          tunnel: [w1557 w1558 w1559 w1560 w1561 w1562 w1563] -> w1452
          tunnel: w1419 -> [_ _ _ _ w1561 _ _]
          tunnel: w1418 -> [_ _ _ _ _ w1562 _]
          tunnel: w1417 -> [_ _ _ _ _ _ w1563]
          frame 0, Default {
          }
          frame 1 {
          }
          frame 2 {
          }
          frame 3 {
          }
          frame 4 {
          }
          frame 5 {
          }
          frame 6 {
          }
        }
        n812 = Equal?(x=w1415, y="W单环Ca") -> (x = y?=w1435:bool)
        n813 = Equal?(x=w1415, y="W单环Cb") -> (x = y?=w1433:bool)
        n814 = Equal?(x=w1415, y="W单环Cc") -> (x = y?=w1434:bool)
        n815 = Equal?(x=w1415, y="W单环Aa") -> (x = y?=w1461:bool)
        n816 = Equal?(x=w1415, y="W单环Ab") -> (x = y?=w1462:bool)
        n817 = Equal?(x=w1415, y="W单环Ac") -> (x = y?=w1448:bool)
        n818 = Equal?(x=w1415, y="W单环Ba") -> (x = y?=w1455:bool)
        n819 = Equal?(x=w1415, y="W单环Bb") -> (x = y?=w1459:bool)
        n820 = Equal?(x=w1415, y="W单环Bc") -> (x = y?=w1457:bool)
        n821 = case shown="True" w1461 {
          tunnel: w1445 -> [w1631 _]
          tunnel: w1416 -> [w1628 _]
          tunnel: w1414 -> [w1627 _]
          frame True {
            n822 = call "绘图-分段颜色-单环.vi"("分段颜色"=w1628, "基准索引"=w1627, "光谱值"=w1631, "清空"="R单环Aa") -> ("数组"=→"F单环Aa":dbl[][])  [unwired: 7 in]
            n823 = case shown="True" "R单环Aa" {
              selector: "R单环Aa" -> [_ w1633]
              frame False {
              }
              frame True {
                n824 = Not(x=w1633) -> (.not. x?=w1632:bool)
                n825 = local write "R单环Aa"(w1632) -> ()
              }
            }
            "N单环Aa" <- w1631
          }
          frame False {
          }
        }
        n826 = case shown="True" w1434 {
          tunnel: w1438 -> [w1498 _]
          tunnel: w1414 -> [w1487 _]
          frame True {
            n827 = feedback #5() -> (w1490:dbl[])  [unwired: 1 in]
            n828 = Select(t=dbl[] [], s="R单环Cc", f=w1490) -> (s? t:f=w1489:dbl[])
            n829 = Build Array (concatenate)(w1489, w1498) -> (w1493:dbl[])
            n830 = feedback-in #5(w1493) -> ()
            n831 = Index Array(array=w1493, index=w1487) -> (element=w1494:dbl)
            n832 = Divide(x=w1494, y=w1493) -> (x/y=w1496:dbl[])
            n833 = Greater Than 0?(x=w1487) -> (x > 0?=w1497:bool)
            n834 = Natural Logarithm(1:w1496) -> (0:w1495:dbl[])
            n835 = Select(t=w1495, s=w1497, f=w1493) -> (s? t:f=→"F单环Cc":dbl[])
            n836 = case shown="True" "R单环Cc" {
              selector: "R单环Cc" -> [_ w1500]
              frame False {
              }
              frame True {
                n837 = Not(x=w1500) -> (.not. x?=w1499:bool)
                n838 = local write "R单环Cc"(w1499) -> ()
              }
            }
            "N单环Cc" <- w1498
          }
          frame False {
          }
        }
        n839 = case shown="True" w1462 {
          tunnel: w1446 -> [w1624 _]
          tunnel: w1414 -> [w1613 _]
          frame True {
            n840 = feedback #6() -> (w1616:dbl[])  [unwired: 1 in]
            n841 = Select(t=dbl[] [], s="R单环Ab", f=w1616) -> (s? t:f=w1615:dbl[])
            n842 = Build Array (concatenate)(w1615, w1624) -> (w1619:dbl[])
            n843 = feedback-in #6(w1619) -> ()
            n844 = Index Array(array=w1619, index=w1613) -> (element=w1620:dbl)
            n845 = Divide(x=w1620, y=w1619) -> (x/y=w1622:dbl[])
            n846 = Greater Than 0?(x=w1613) -> (x > 0?=w1623:bool)
            n847 = Natural Logarithm(1:w1622) -> (0:w1621:dbl[])
            n848 = Select(t=w1621, s=w1623, f=w1619) -> (s? t:f=→"F单环Ab":dbl[])
            n849 = case shown="True" "R单环Ab" {
              selector: "R单环Ab" -> [_ w1626]
              frame False {
              }
              frame True {
                n850 = Not(x=w1626) -> (.not. x?=w1625:bool)
                n851 = local write "R单环Ab"(w1625) -> ()
              }
            }
            "N单环Ab" <- w1624
          }
          frame False {
          }
        }
        n852 = case shown="True" w1457 {
          tunnel: w1452 -> [w1589 _]
          tunnel: w1414 -> [w1578 _]
          frame True {
            n853 = feedback #7() -> (w1581:dbl[])  [unwired: 1 in]
            n854 = Select(t=dbl[] [], s="R单环Bc", f=w1581) -> (s? t:f=w1580:dbl[])
            n855 = Build Array (concatenate)(w1580, w1589) -> (w1584:dbl[])
            n856 = feedback-in #7(w1584) -> ()
            n857 = Index Array(array=w1584, index=w1578) -> (element=w1583:dbl)
            n858 = Divide(x=w1583, y=w1584) -> (x/y=w1587:dbl[])
            n859 = Greater Than 0?(x=w1578) -> (x > 0?=w1588:bool)
            n860 = Natural Logarithm(1:w1587) -> (0:w1586:dbl[])
            n861 = Select(t=w1586, s=w1588, f=w1584) -> (s? t:f=→"F单环Bc":dbl[])
            n862 = case shown="True" "R单环Bc" {
              selector: "R单环Bc" -> [_ w1591]
              frame False {
              }
              frame True {
                n863 = Not(x=w1591) -> (.not. x?=w1590:bool)
                n864 = local write "R单环Bc"(w1590) -> ()
              }
            }
            "N单环Bc" <- w1589
          }
          frame False {
          }
        }
        n865 = case shown="True" w1433 {
          tunnel: w1437 -> [w1512 _]
          tunnel: w1414 -> [w1501 _]
          frame True {
            n866 = feedback #8() -> (w1504:dbl[])  [unwired: 1 in]
            n867 = Select(t=dbl[] [], s="R单环Cb", f=w1504) -> (s? t:f=w1503:dbl[])
            n868 = Build Array (concatenate)(w1503, w1512) -> (w1506:dbl[])
            n869 = feedback-in #8(w1506) -> ()
            n870 = Index Array(array=w1506, index=w1501) -> (element=w1507:dbl)
            n871 = Divide(x=w1507, y=w1506) -> (x/y=w1510:dbl[])
            n872 = Greater Than 0?(x=w1501) -> (x > 0?=w1511:bool)
            n873 = Natural Logarithm(1:w1510) -> (0:w1509:dbl[])
            n874 = Select(t=w1509, s=w1511, f=w1506) -> (s? t:f=→"F单环Cb":dbl[])
            n875 = case shown="True" "R单环Cb" {
              selector: "R单环Cb" -> [_ w1514]
              frame False {
              }
              frame True {
                n876 = Not(x=w1514) -> (.not. x?=w1513:bool)
                n877 = local write "R单环Cb"(w1513) -> ()
              }
            }
            "N单环Cb" <- w1512
          }
          frame False {
          }
        }
        n878 = case shown="True" w1448 {
          tunnel: w1447 -> [w1554 _]
          tunnel: w1414 -> [w1543 _]
          frame True {
            n879 = feedback #9() -> (w1546:dbl[])  [unwired: 1 in]
            n880 = Select(t=dbl[] [], s="R单环Ac", f=w1546) -> (s? t:f=w1545:dbl[])
            n881 = Build Array (concatenate)(w1545, w1554) -> (w1549:dbl[])
            n882 = feedback-in #9(w1549) -> ()
            n883 = Index Array(array=w1549, index=w1543) -> (element=w1550:dbl)
            n884 = Divide(x=w1550, y=w1549) -> (x/y=w1552:dbl[])
            n885 = Greater Than 0?(x=w1543) -> (x > 0?=w1553:bool)
            n886 = Natural Logarithm(1:w1552) -> (0:w1551:dbl[])
            n887 = Select(t=w1551, s=w1553, f=w1549) -> (s? t:f=→"F单环Ac":dbl[])
            n888 = case shown="True" "R单环Ac" {
              selector: "R单环Ac" -> [_ w1556]
              frame False {
              }
              frame True {
                n889 = Not(x=w1556) -> (.not. x?=w1555:bool)
                n890 = local write "R单环Ac"(w1555) -> ()
              }
            }
            "N单环Ac" <- w1554
          }
          frame False {
          }
        }
        n891 = case shown="True" w1459 {
          tunnel: w1453 -> [w1603 _]
          tunnel: w1414 -> [w1592 _]
          frame True {
            n892 = feedback #10() -> (w1594:dbl[])  [unwired: 1 in]
            n893 = Select(t=dbl[] [], s="R单环Bb", f=w1594) -> (s? t:f=w1595:dbl[])
            n894 = Build Array (concatenate)(w1595, w1603) -> (w1599:dbl[])
            n895 = feedback-in #10(w1599) -> ()
            n896 = Index Array(array=w1599, index=w1592) -> (element=w1598:dbl)
            n897 = Divide(x=w1598, y=w1599) -> (x/y=w1601:dbl[])
            n898 = Greater Than 0?(x=w1592) -> (x > 0?=w1602:bool)
            n899 = Natural Logarithm(1:w1601) -> (0:w1600:dbl[])
            n900 = Select(t=w1600, s=w1602, f=w1599) -> (s? t:f=→"F单环Bb":dbl[])
            n901 = case shown="True" "R单环Bb" {
              selector: "R单环Bb" -> [_ w1605]
              frame False {
              }
              frame True {
                n902 = Not(x=w1605) -> (.not. x?=w1604:bool)
                n903 = local write "R单环Bb"(w1604) -> ()
              }
            }
            "N单环Bb" <- w1603
          }
          frame False {
          }
        }
        n904 = case shown="True" w1435 {
          tunnel: w1436 -> [w1517 _]
          tunnel: w1416 -> [w1519 _]
          tunnel: w1414 -> [w1515 _]
          frame True {
            n905 = call "绘图-分段颜色-单环.vi"("分段颜色"=w1519, "基准索引"=w1515, "光谱值"=w1517, "清空"="R单环Ca") -> ("数组"=→"F单环Ca":dbl[][])  [unwired: 7 in]
            n906 = case shown="True" "R单环Ca" {
              selector: "R单环Ca" -> [_ w1521]
              frame False {
              }
              frame True {
                n907 = Not(x=w1521) -> (.not. x?=w1520:bool)
                n908 = local write "R单环Ca"(w1520) -> ()
              }
            }
            "N单环Ca" <- w1517
          }
          frame False {
          }
        }
        n909 = case shown="True" w1455 {
          tunnel: w1454 -> [w1610 _]
          tunnel: w1416 -> [w1608 _]
          tunnel: w1414 -> [w1606 _]
          frame True {
            n910 = call "绘图-分段颜色-单环.vi"("分段颜色"=w1608, "基准索引"=w1606, "光谱值"=w1610, "清空"="R单环Ba") -> ("数组"=→"F单环Ba":dbl[][])  [unwired: 7 in]
            n911 = case shown="True" "R单环Ba" {
              selector: "R单环Ba" -> [_ w1612]
              frame False {
              }
              frame True {
                n912 = Not(x=w1612) -> (.not. x?=w1611:bool)
                n913 = local write "R单环Ba"(w1611) -> ()
              }
            }
            "N单环Ba" <- w1610
          }
          frame False {
          }
        }
        n914 = call <vilib>:"Add State(s) to Queue__JKI_lib_State_Machine.vi"("State(s) in (\"\")"=w1463) -> ("States Out"=w1464:string)  [unwired: 14 in]
      }
      frame "UI: Update Graph_Diff_LT1" {
        # "长期-差分1"
        n915 = Unbundle By Name(w1643) -> ("Time and Data.当前运行信息.当前索引子集"=w1645:i8[], "Indicators.图表相关.分段颜色"=w1644:enum32{"蓝色", "红色"}, "Time and Data.Data"=w1719:dbl[], "Sample Settings.校准.温度校准值"=w1646:dbl[], "Indicators.图表相关.基准索引"=w1634:i32)
        n916 = Index Array(array=w1645) -> (element=w1635:i8)  [unwired: 1 in]
        n917 = Index Array(array=w1719) -> (element #1=w1642:dbl, element #2=w1641:dbl, element #3=w1640:dbl, element #4=w1639:dbl, element #5=w1638:dbl, element #6=w1637:dbl, element #7=w1636:dbl)  [unwired: 7 in]
        n918 = case shown="20" "差分Ab" {
          tunnel: w1642 -> [w2018 w2020 w2022 w2024 _ _ _ _ _ _ w2038 w2040 _ _ _ _ _ _ _ _ _]
          tunnel: w1641 -> [w2017 _ _ _ w2026 w2028 w2030 _ _ _ _ _ w2042 w2044 _ _ _ _ _ _ _]
          tunnel: w1640 -> [_ w2019 _ _ w2025 _ _ w2032 w2034 _ _ _ _ _ w2046 w2048 _ _ _ _ _]
          tunnel: w1639 -> [_ _ w2021 _ _ w2027 _ w2031 _ w2036 _ _ _ _ _ _ w2050 w2052 _ _ _]
          tunnel: [w2018 w2020 w2022 w2024 w2026 w2028 w2030 w2032 w2034 w2036 w2038 w2040 w2042 w2044 w2046 w2048 w2050 w2052 w2054 w2056 w2058] -> w1671
          tunnel: [w2017 w2019 w2021 w2023 w2025 w2027 w2029 w2031 w2033 w2035 w2037 w2039 w2041 w2043 w2045 w2047 w2049 w2051 w2053 w2055 w2057] -> w1670
          tunnel: w1638 -> [_ _ _ w2023 _ _ w2029 _ w2033 w2035 _ _ _ _ _ _ _ _ w2054 w2056 _]
          tunnel: w1637 -> [_ _ _ _ _ _ _ _ _ _ w2037 _ w2041 _ w2045 _ w2049 _ w2053 _ w2058]
          tunnel: w1636 -> [_ _ _ _ _ _ _ _ _ _ _ w2039 _ w2043 _ w2047 _ w2051 _ w2055 w2057]
          frame 0, Default {
          }
          frame 1 {
          }
          frame 2 {
          }
          frame 3 {
          }
          frame 4 {
          }
          frame 5 {
          }
          frame 6 {
          }
          frame 7 {
          }
          frame 8 {
          }
          frame 9 {
          }
          frame 10 {
          }
          frame 11 {
          }
          frame 12 {
          }
          frame 13 {
          }
          frame 14 {
          }
          frame 15 {
          }
          frame 16 {
          }
          frame 17 {
          }
          frame 18 {
          }
          frame 19 {
          }
          frame 20 {
          }
        }
        n919 = case shown="20" "差分Ba" {
          tunnel: w1642 -> [w1934 w1936 w1938 w1940 _ _ _ _ _ _ w1954 w1956 _ _ _ _ _ _ _ _ _]
          tunnel: w1641 -> [w1933 _ _ _ w1942 w1944 w1946 _ _ _ _ _ w1958 w1960 _ _ _ _ _ _ _]
          tunnel: w1640 -> [_ w1935 _ _ w1941 _ _ w1948 w1950 _ _ _ _ _ w1962 w1964 _ _ _ _ _]
          tunnel: w1639 -> [_ _ w1937 _ _ w1943 _ w1947 _ w1952 _ _ _ _ _ _ w1966 w1968 _ _ _]
          tunnel: [w1934 w1936 w1938 w1940 w1942 w1944 w1946 w1948 w1950 w1952 w1954 w1956 w1958 w1960 w1962 w1964 w1966 w1968 w1970 w1972 w1974] -> w1665
          tunnel: [w1933 w1935 w1937 w1939 w1941 w1943 w1945 w1947 w1949 w1951 w1953 w1955 w1957 w1959 w1961 w1963 w1965 w1967 w1969 w1971 w1973] -> w1664
          tunnel: w1638 -> [_ _ _ w1939 _ _ w1945 _ w1949 w1951 _ _ _ _ _ _ _ _ w1970 w1972 _]
          tunnel: w1637 -> [_ _ _ _ _ _ _ _ _ _ w1953 _ w1957 _ w1961 _ w1965 _ w1969 _ w1974]
          tunnel: w1636 -> [_ _ _ _ _ _ _ _ _ _ _ w1955 _ w1959 _ w1963 _ w1967 _ w1971 w1973]
          frame 0, Default {
          }
          frame 1 {
          }
          frame 2 {
          }
          frame 3 {
          }
          frame 4 {
          }
          frame 5 {
          }
          frame 6 {
          }
          frame 7 {
          }
          frame 8 {
          }
          frame 9 {
          }
          frame 10 {
          }
          frame 11 {
          }
          frame 12 {
          }
          frame 13 {
          }
          frame 14 {
          }
          frame 15 {
          }
          frame 16 {
          }
          frame 17 {
          }
          frame 18 {
          }
          frame 19 {
          }
          frame 20 {
          }
        }
        n920 = case shown="20" "差分Bb" {
          tunnel: w1642 -> [w1892 w1894 w1896 w1898 _ _ _ _ _ _ w1912 w1914 _ _ _ _ _ _ _ _ _]
          tunnel: w1641 -> [w1891 _ _ _ w1900 w1902 w1904 _ _ _ _ _ w1916 w1918 _ _ _ _ _ _ _]
          tunnel: w1640 -> [_ w1893 _ _ w1899 _ _ w1906 w1908 _ _ _ _ _ w1920 w1922 _ _ _ _ _]
          tunnel: w1639 -> [_ _ w1895 _ _ w1901 _ w1905 _ w1910 _ _ _ _ _ _ w1924 w1926 _ _ _]
          tunnel: [w1892 w1894 w1896 w1898 w1900 w1902 w1904 w1906 w1908 w1910 w1912 w1914 w1916 w1918 w1920 w1922 w1924 w1926 w1928 w1930 w1932] -> w1661
          tunnel: [w1891 w1893 w1895 w1897 w1899 w1901 w1903 w1905 w1907 w1909 w1911 w1913 w1915 w1917 w1919 w1921 w1923 w1925 w1927 w1929 w1931] -> w1660
          tunnel: w1638 -> [_ _ _ w1897 _ _ w1903 _ w1907 w1909 _ _ _ _ _ _ _ _ w1928 w1930 _]
          tunnel: w1637 -> [_ _ _ _ _ _ _ _ _ _ w1911 _ w1915 _ w1919 _ w1923 _ w1927 _ w1932]
          tunnel: w1636 -> [_ _ _ _ _ _ _ _ _ _ _ w1913 _ w1917 _ w1921 _ w1925 _ w1929 w1931]
          frame 0, Default {
          }
          frame 1 {
          }
          frame 2 {
          }
          frame 3 {
          }
          frame 4 {
          }
          frame 5 {
          }
          frame 6 {
          }
          frame 7 {
          }
          frame 8 {
          }
          frame 9 {
          }
          frame 10 {
          }
          frame 11 {
          }
          frame 12 {
          }
          frame 13 {
          }
          frame 14 {
          }
          frame 15 {
          }
          frame 16 {
          }
          frame 17 {
          }
          frame 18 {
          }
          frame 19 {
          }
          frame 20 {
          }
        }
        n921 = case shown="20" "差分Ca" {
          tunnel: w1642 -> [w1850 w1852 w1854 w1856 _ _ _ _ _ _ w1870 w1872 _ _ _ _ _ _ _ _ _]
          tunnel: w1641 -> [w1849 _ _ _ w1858 w1860 w1862 _ _ _ _ _ w1874 w1876 _ _ _ _ _ _ _]
          tunnel: w1640 -> [_ w1851 _ _ w1857 _ _ w1864 w1866 _ _ _ _ _ w1878 w1880 _ _ _ _ _]
          tunnel: w1639 -> [_ _ w1853 _ _ w1859 _ w1863 _ w1868 _ _ _ _ _ _ w1882 w1884 _ _ _]
          tunnel: [w1850 w1852 w1854 w1856 w1858 w1860 w1862 w1864 w1866 w1868 w1870 w1872 w1874 w1876 w1878 w1880 w1882 w1884 w1886 w1888 w1890] -> w1658
          tunnel: [w1849 w1851 w1853 w1855 w1857 w1859 w1861 w1863 w1865 w1867 w1869 w1871 w1873 w1875 w1877 w1879 w1881 w1883 w1885 w1887 w1889] -> w1657
          tunnel: w1638 -> [_ _ _ w1855 _ _ w1861 _ w1865 w1867 _ _ _ _ _ _ _ _ w1886 w1888 _]
          tunnel: w1637 -> [_ _ _ _ _ _ _ _ _ _ w1869 _ w1873 _ w1877 _ w1881 _ w1885 _ w1890]
          tunnel: w1636 -> [_ _ _ _ _ _ _ _ _ _ _ w1871 _ w1875 _ w1879 _ w1883 _ w1887 w1889]
          frame 0, Default {
          }
          frame 1 {
          }
          frame 2 {
          }
          frame 3 {
          }
          frame 4 {
          }
          frame 5 {
          }
          frame 6 {
          }
          frame 7 {
          }
          frame 8 {
          }
          frame 9 {
          }
          frame 10 {
          }
          frame 11 {
          }
          frame 12 {
          }
          frame 13 {
          }
          frame 14 {
          }
          frame 15 {
          }
          frame 16 {
          }
          frame 17 {
          }
          frame 18 {
          }
          frame 19 {
          }
          frame 20 {
          }
        }
        n922 = case shown="20" "差分Cb" {
          tunnel: w1642 -> [w1766 w1768 w1770 w1772 _ _ _ _ _ _ w1786 w1788 _ _ _ _ _ _ _ _ _]
          tunnel: w1641 -> [w1765 _ _ _ w1774 w1776 w1778 _ _ _ _ _ w1790 w1792 _ _ _ _ _ _ _]
          tunnel: w1640 -> [_ w1767 _ _ w1773 _ _ w1780 w1782 _ _ _ _ _ w1794 w1796 _ _ _ _ _]
          tunnel: w1639 -> [_ _ w1769 _ _ w1775 _ w1779 _ w1784 _ _ _ _ _ _ w1798 w1800 _ _ _]
          tunnel: [w1766 w1768 w1770 w1772 w1774 w1776 w1778 w1780 w1782 w1784 w1786 w1788 w1790 w1792 w1794 w1796 w1798 w1800 w1802 w1804 w1806] -> w1652
          tunnel: [w1765 w1767 w1769 w1771 w1773 w1775 w1777 w1779 w1781 w1783 w1785 w1787 w1789 w1791 w1793 w1795 w1797 w1799 w1801 w1803 w1805] -> w1651
          tunnel: w1638 -> [_ _ _ w1771 _ _ w1777 _ w1781 w1783 _ _ _ _ _ _ _ _ w1802 w1804 _]
          tunnel: w1637 -> [_ _ _ _ _ _ _ _ _ _ w1785 _ w1789 _ w1793 _ w1797 _ w1801 _ w1806]
          tunnel: w1636 -> [_ _ _ _ _ _ _ _ _ _ _ w1787 _ w1791 _ w1795 _ w1799 _ w1803 w1805]
          frame 0, Default {
          }
          frame 1 {
          }
          frame 2 {
          }
          frame 3 {
          }
          frame 4 {
          }
          frame 5 {
          }
          frame 6 {
          }
          frame 7 {
          }
          frame 8 {
          }
          frame 9 {
          }
          frame 10 {
          }
          frame 11 {
          }
          frame 12 {
          }
          frame 13 {
          }
          frame 14 {
          }
          frame 15 {
          }
          frame 16 {
          }
          frame 17 {
          }
          frame 18 {
          }
          frame 19 {
          }
          frame 20 {
          }
        }
        n923 = case shown="20" "差分Cc" {
          tunnel: w1642 -> [w1724 w1726 w1728 w1730 _ _ _ _ _ _ w1744 w1746 _ _ _ _ _ _ _ _ _]
          tunnel: w1641 -> [w1723 _ _ _ w1732 w1734 w1736 _ _ _ _ _ w1748 w1750 _ _ _ _ _ _ _]
          tunnel: w1640 -> [_ w1725 _ _ w1731 _ _ w1738 w1740 _ _ _ _ _ w1752 w1754 _ _ _ _ _]
          tunnel: w1639 -> [_ _ w1727 _ _ w1733 _ w1737 _ w1742 _ _ _ _ _ _ w1756 w1758 _ _ _]
          tunnel: [w1724 w1726 w1728 w1730 w1732 w1734 w1736 w1738 w1740 w1742 w1744 w1746 w1748 w1750 w1752 w1754 w1756 w1758 w1760 w1762 w1764] -> w1649
          tunnel: [w1723 w1725 w1727 w1729 w1731 w1733 w1735 w1737 w1739 w1741 w1743 w1745 w1747 w1749 w1751 w1753 w1755 w1757 w1759 w1761 w1763] -> w1648
          tunnel: w1638 -> [_ _ _ w1729 _ _ w1735 _ w1739 w1741 _ _ _ _ _ _ _ _ w1760 w1762 _]
          tunnel: w1637 -> [_ _ _ _ _ _ _ _ _ _ w1743 _ w1747 _ w1751 _ w1755 _ w1759 _ w1764]
          tunnel: w1636 -> [_ _ _ _ _ _ _ _ _ _ _ w1745 _ w1749 _ w1753 _ w1757 _ w1761 w1763]
          frame 0, Default {
          }
          frame 1 {
          }
          frame 2 {
          }
          frame 3 {
          }
          frame 4 {
          }
          frame 5 {
          }
          frame 6 {
          }
          frame 7 {
          }
          frame 8 {
          }
          frame 9 {
          }
          frame 10 {
          }
          frame 11 {
          }
          frame 12 {
          }
          frame 13 {
          }
          frame 14 {
          }
          frame 15 {
          }
          frame 16 {
          }
          frame 17 {
          }
          frame 18 {
          }
          frame 19 {
          }
          frame 20 {
          }
        }
        n924 = case shown="0, 默认" "差分Aa" {
          tunnel: w1642 -> [w2070 w2072 w2074 w2076 _ _ _ _ _ _ w2090 w2092 _ _ _ _ _ _ _ _ _]
          tunnel: w1641 -> [w2069 _ _ _ w2078 w2080 w2082 _ _ _ _ _ w2094 w2096 _ _ _ _ _ _ _]
          tunnel: w1640 -> [_ w2071 _ _ w2077 _ _ w2084 w2086 _ _ _ _ _ w2098 w2100 _ _ _ _ _]
          tunnel: w1639 -> [_ _ w2073 _ _ w2079 _ w2083 _ w2088 _ _ _ _ _ _ w2102 w2104 _ _ _]
          tunnel: [w2070 w2072 w2074 w2076 w2078 w2080 w2082 w2084 w2086 w2088 w2090 w2092 w2094 w2096 w2098 w2100 w2102 w2104 w2106 w2108 w2110] -> w1701
          tunnel: [w2069 w2071 w2073 w2075 w2077 w2079 w2081 w2083 w2085 w2087 w2089 w2091 w2093 w2095 w2097 w2099 w2101 w2103 w2105 w2107 w2109] -> w1702
          tunnel: w1638 -> [_ _ _ w2075 _ _ w2081 _ w2085 w2087 _ _ _ _ _ _ _ _ w2106 w2108 _]
          tunnel: w1637 -> [_ _ _ _ _ _ _ _ _ _ w2089 _ w2093 _ w2097 _ w2101 _ w2105 _ w2110]
          tunnel: w1636 -> [_ _ _ _ _ _ _ _ _ _ _ w2091 _ w2095 _ w2099 _ w2103 _ w2107 w2109]
          frame 0, Default {
          }
          frame 1 {
          }
          frame 2 {
          }
          frame 3 {
          }
          frame 4 {
          }
          frame 5 {
          }
          frame 6 {
          }
          frame 7 {
          }
          frame 8 {
          }
          frame 9 {
          }
          frame 10 {
          }
          frame 11 {
          }
          frame 12 {
          }
          frame 13 {
          }
          frame 14 {
          }
          frame 15 {
          }
          frame 16 {
          }
          frame 17 {
          }
          frame 18 {
          }
          frame 19 {
          }
          frame 20 {
          }
        }
        n925 = case shown="20" "差分Ac" {
          tunnel: w1642 -> [w1976 w1978 w1980 w1982 _ _ _ _ _ _ w1996 w1998 _ _ _ _ _ _ _ _ _]
          tunnel: w1641 -> [w1975 _ _ _ w1984 w1986 w1988 _ _ _ _ _ w2000 w2002 _ _ _ _ _ _ _]
          tunnel: w1640 -> [_ w1977 _ _ w1983 _ _ w1990 w1992 _ _ _ _ _ w2004 w2006 _ _ _ _ _]
          tunnel: w1639 -> [_ _ w1979 _ _ w1985 _ w1989 _ w1994 _ _ _ _ _ _ w2008 w2010 _ _ _]
          tunnel: [w1976 w1978 w1980 w1982 w1984 w1986 w1988 w1990 w1992 w1994 w1996 w1998 w2000 w2002 w2004 w2006 w2008 w2010 w2012 w2014 w2016] -> w1667
          tunnel: [w1975 w1977 w1979 w1981 w1983 w1985 w1987 w1989 w1991 w1993 w1995 w1997 w1999 w2001 w2003 w2005 w2007 w2009 w2011 w2013 w2015] -> w1666
          tunnel: w1638 -> [_ _ _ w1981 _ _ w1987 _ w1991 w1993 _ _ _ _ _ _ _ _ w2012 w2014 _]
          tunnel: w1637 -> [_ _ _ _ _ _ _ _ _ _ w1995 _ w1999 _ w2003 _ w2007 _ w2011 _ w2016]
          tunnel: w1636 -> [_ _ _ _ _ _ _ _ _ _ _ w1997 _ w2001 _ w2005 _ w2009 _ w2013 w2015]
          frame 0, Default {
          }
          frame 1 {
          }
          frame 2 {
          }
          frame 3 {
          }
          frame 4 {
          }
          frame 5 {
          }
          frame 6 {
          }
          frame 7 {
          }
          frame 8 {
          }
          frame 9 {
          }
          frame 10 {
          }
          frame 11 {
          }
          frame 12 {
          }
          frame 13 {
          }
          frame 14 {
          }
          frame 15 {
          }
          frame 16 {
          }
          frame 17 {
          }
          frame 18 {
          }
          frame 19 {
          }
          frame 20 {
          }
        }
        n926 = case shown="20" "差分Bc" {
          tunnel: w1642 -> [w1808 w1810 w1812 w1814 _ _ _ _ _ _ w1828 w1830 _ _ _ _ _ _ _ _ _]
          tunnel: w1641 -> [w1807 _ _ _ w1816 w1818 w1820 _ _ _ _ _ w1832 w1834 _ _ _ _ _ _ _]
          tunnel: w1640 -> [_ w1809 _ _ w1815 _ _ w1822 w1824 _ _ _ _ _ w1836 w1838 _ _ _ _ _]
          tunnel: w1639 -> [_ _ w1811 _ _ w1817 _ w1821 _ w1826 _ _ _ _ _ _ w1840 w1842 _ _ _]
          tunnel: [w1808 w1810 w1812 w1814 w1816 w1818 w1820 w1822 w1824 w1826 w1828 w1830 w1832 w1834 w1836 w1838 w1840 w1842 w1844 w1846 w1848] -> w1655
          tunnel: [w1807 w1809 w1811 w1813 w1815 w1817 w1819 w1821 w1823 w1825 w1827 w1829 w1831 w1833 w1835 w1837 w1839 w1841 w1843 w1845 w1847] -> w1654
          tunnel: w1638 -> [_ _ _ w1813 _ _ w1819 _ w1823 w1825 _ _ _ _ _ _ _ _ w1844 w1846 _]
          tunnel: w1637 -> [_ _ _ _ _ _ _ _ _ _ w1827 _ w1831 _ w1835 _ w1839 _ w1843 _ w1848]
          tunnel: w1636 -> [_ _ _ _ _ _ _ _ _ _ _ w1829 _ w1833 _ w1837 _ w1841 _ w1845 w1847]
          frame 0, Default {
          }
          frame 1 {
          }
          frame 2 {
          }
          frame 3 {
          }
          frame 4 {
          }
          frame 5 {
          }
          frame 6 {
          }
          frame 7 {
          }
          frame 8 {
          }
          frame 9 {
          }
          frame 10 {
          }
          frame 11 {
          }
          frame 12 {
          }
          frame 13 {
          }
          frame 14 {
          }
          frame 15 {
          }
          frame 16 {
          }
          frame 17 {
          }
          frame 18 {
          }
          frame 19 {
          }
          frame 20 {
          }
        }
        n927 = xnode "公式 Cb"("X1"=w1652, "X2"=w1651) -> ("结果"=w1694:dbl)  [unwired: 1 in, 1 out]
        n928 = xnode "公式 Cc"("X1"=w1649, "X2"=w1648) -> ("结果"=w1697:dbl)  [unwired: 1 in, 1 out]
        n929 = xnode "公式 Aa"("X1"=w1701, "X2"=w1702) -> ("结果"=w1673:dbl)  [unwired: 1 in, 1 out]
        n930 = xnode "公式 Ab"("X1"=w1671, "X2"=w1670) -> ("结果"=w1676:dbl)  [unwired: 1 in, 1 out]
        n931 = xnode "公式 Ba"("X1"=w1665, "X2"=w1664) -> ("结果"=w1681:dbl)  [unwired: 1 in, 1 out]
        n932 = xnode "公式 Bb"("X1"=w1661, "X2"=w1660) -> ("结果"=w1685:dbl)  [unwired: 1 in, 1 out]
        n933 = xnode "公式 Ca"("X1"=w1658, "X2"=w1657) -> ("结果"=w1691:dbl)  [unwired: 1 in, 1 out]
        n934 = xnode "公式 Ac"("X1"=w1667, "X2"=w1666) -> ("结果"=w1679:dbl)  [unwired: 1 in, 1 out]
        n935 = xnode "公式 Bc"("X1"=w1655, "X2"=w1654) -> ("结果"=w1688:dbl)  [unwired: 1 in, 1 out]
        n936 = Index Array(array=w1646, index="差分Ba") -> (element=w1682:dbl)
        n937 = Index Array(array=w1646, index="差分Cb") -> (element=w1693:dbl)
        n938 = Index Array(array=w1646, index="差分Ab") -> (element=w1675:dbl)
        n939 = Index Array(array=w1646, index="差分Ac") -> (element=w1678:dbl)
        n940 = Index Array(array=w1646, index="差分Bc") -> (element=w1687:dbl)
        n941 = Index Array(array=w1646, index="差分Aa") -> (element=w1672:dbl)
        n942 = Index Array(array=w1646, index="差分Bb") -> (element=w1684:dbl)
        n943 = Index Array(array=w1646, index="差分Ca") -> (element=w1690:dbl)
        n944 = Index Array(array=w1646, index="差分Cc") -> (element=w1696:dbl)
        n945 = Subtract(x=w1679, y=w1678) -> (x-y=w1677:dbl)
        n946 = Subtract(x=w1681, y=w1682) -> (x-y=w1680:dbl)
        n947 = Subtract(x=w1676, y=w1675) -> (x-y=w1674:dbl)
        n948 = Subtract(x=w1673, y=w1672) -> (x-y=w1647:dbl)
        n949 = Subtract(x=w1685, y=w1684) -> (x-y=w1683:dbl)
        n950 = Subtract(x=w1688, y=w1687) -> (x-y=w1686:dbl)
        n951 = Subtract(x=w1694, y=w1693) -> (x-y=w1692:dbl)
        n952 = Subtract(x=w1691, y=w1690) -> (x-y=w1689:dbl)
        n953 = Subtract(x=w1697, y=w1696) -> (x-y=w1695:dbl)
        n954 = Equal?(x=w1635, y="W差分Aa") -> (x = y?=w1700:bool)
        n955 = Equal?(x=w1635, y="W差分Ab") -> (x = y?=w1717:bool)
        n956 = Equal?(x=w1635, y="W差分Ac") -> (x = y?=w1715:bool)
        n957 = Equal?(x=w1635, y="W差分Ba") -> (x = y?=w1713:bool)
        n958 = Equal?(x=w1635, y="W差分Bb") -> (x = y?=w1707:bool)
        n959 = Equal?(x=w1635, y="W差分Bc") -> (x = y?=w1703:bool)
        n960 = Equal?(x=w1635, y="W差分Ca") -> (x = y?=w1709:bool)
        n961 = Equal?(x=w1635, y="W差分Cb") -> (x = y?=w1711:bool)
        n962 = Equal?(x=w1635, y="W差分Cc") -> (x = y?=w1705:bool)
        n963 = case shown="True" w1709 {
          tunnel: w1689 -> [w2228 _]
          tunnel: w1644 -> [w2226 _]
          tunnel: w1634 -> [w2224 _]
          frame True {
            n964 = Build Array(w2228) -> (w2225:dbl[])
            n965 = call "绘图-分段颜色-差分.vi"("分段颜色"=w2226, "基准索引"=w2224, "光谱值"=w2225, "清空"="R差分Ca") -> ("数组"=→"F差分Ca":dbl[][])  [unwired: 7 in]
            n966 = case shown="True" "R差分Ca" {
              selector: "R差分Ca" -> [_ w2231]
              frame False {
              }
              frame True {
                n967 = Not(x=w2231) -> (.not. x?=w2230:bool)
                n968 = local write "R差分Ca"(w2230) -> ()
              }
            }
            "N差分Ca" <- w2228
          }
          frame False {
          }
        }
        n969 = case shown="True" w1717 {
          tunnel: w1674 -> [w2268 _]
          tunnel: w1634 -> [w2262 _]
          frame True {
            n970 = feedback #11() -> (w2265:dbl[])  [unwired: 1 in]
            n971 = Select(t=dbl[] [], s="R差分Ab", f=w2265) -> (s? t:f=w2266:dbl[])
            n972 = Build Array (concatenate)(w2266, w2268) -> (w2269:dbl[])
            n973 = feedback-in #11(w2269) -> ()
            n974 = Index Array(array=w2269, index=w2262) -> (element=w2270:dbl)
            n975 = Subtract(x=w2269, y=w2270) -> (x-y=→"F差分Ab":dbl[])
            n976 = case shown="True" "R差分Ab" {
              selector: "R差分Ab" -> [_ w2272]
              frame False {
              }
              frame True {
                n977 = Not(x=w2272) -> (.not. x?=w2271:bool)
                n978 = local write "R差分Ab"(w2271) -> ()
              }
            }
            "N差分Ab" <- w2268
          }
          frame False {
          }
        }
        n979 = case shown="True" w1703 {
          tunnel: w1686 -> [w2197 _]
          tunnel: w1634 -> [w2191 _]
          frame True {
            n980 = feedback #12() -> (w2194:dbl[])  [unwired: 1 in]
            n981 = Select(t=dbl[] [], s="R差分Bc", f=w2194) -> (s? t:f=w2193:dbl[])
            n982 = Build Array (concatenate)(w2193, w2197) -> (w2199:dbl[])
            n983 = feedback-in #12(w2199) -> ()
            n984 = Index Array(array=w2199, index=w2191) -> (element=w2198:dbl)
            n985 = Subtract(x=w2199, y=w2198) -> (x-y=→"F差分Bc":dbl[])
            n986 = case shown="True" "R差分Bc" {
              selector: "R差分Bc" -> [_ w2201]
              frame False {
              }
              frame True {
                n987 = Not(x=w2201) -> (.not. x?=w2200:bool)
                n988 = local write "R差分Bc"(w2200) -> ()
              }
            }
            "N差分Bc" <- w2197
          }
          frame False {
          }
        }
        n989 = case shown="True" w1705 {
          tunnel: w1695 -> [w2208 _]
          tunnel: w1634 -> [w2202 _]
          frame True {
            n990 = feedback #13() -> (w2205:dbl[])  [unwired: 1 in]
            n991 = Select(t=dbl[] [], s="R差分Cc", f=w2205) -> (s? t:f=w2204:dbl[])
            n992 = Build Array (concatenate)(w2204, w2208) -> (w2209:dbl[])
            n993 = feedback-in #13(w2209) -> ()
            n994 = Index Array(array=w2209, index=w2202) -> (element=w2210:dbl)
            n995 = Subtract(x=w2209, y=w2210) -> (x-y=→"F差分Cc":dbl[])
            n996 = case shown="True" "R差分Cc" {
              selector: "R差分Cc" -> [_ w2212]
              frame False {
              }
              frame True {
                n997 = Not(x=w2212) -> (.not. x?=w2211:bool)
                n998 = local write "R差分Cc"(w2211) -> ()
              }
            }
            "N差分Cc" <- w2208
          }
          frame False {
          }
        }
        n999 = case shown="True" w1715 {
          tunnel: w1677 -> [w2255 _]
          tunnel: w1634 -> [w2251 _]
          frame True {
            n1000 = feedback #14() -> (w2256:dbl[])  [unwired: 1 in]
            n1001 = Select(t=dbl[] [], s="R差分Ac", f=w2256) -> (s? t:f=w2259:dbl[])
            n1002 = Build Array (concatenate)(w2259, w2255) -> (w2254:dbl[])
            n1003 = feedback-in #14(w2254) -> ()
            n1004 = Index Array(array=w2254, index=w2251) -> (element=w2253:dbl)
            n1005 = case shown="True" "R差分Ac" {
              selector: "R差分Ac" -> [_ w2261]
              frame False {
              }
              frame True {
                n1006 = Not(x=w2261) -> (.not. x?=w2260:bool)
                n1007 = local write "R差分Ac"(w2260) -> ()
              }
            }
            n1008 = Subtract(x=w2254, y=w2253) -> (x-y=→"F差分Ac":dbl[])
            "N差分Ac" <- w2255
          }
          frame False {
          }
        }
        n1009 = case shown="True" w1713 {
          tunnel: w1680 -> [w2245 _]
          tunnel: w1644 -> [w2246 _]
          tunnel: w1634 -> [w2243 _]
          frame True {
            n1010 = Build Array(w2245) -> (w2244:dbl[])
            n1011 = call "绘图-分段颜色-差分.vi"("分段颜色"=w2246, "基准索引"=w2243, "光谱值"=w2244, "清空"="R差分Ba") -> ("数组"=→"F差分Ba":dbl[][])  [unwired: 7 in]
            n1012 = case shown="True" "R差分Ba" {
              selector: "R差分Ba" -> [_ w2250]
              frame False {
              }
              frame True {
                n1013 = Not(x=w2250) -> (.not. x?=w2249:bool)
                n1014 = local write "R差分Ba"(w2249) -> ()
              }
            }
            "N差分Ba" <- w2245
          }
          frame False {
          }
        }
        n1015 = case shown="True" w1707 {
          tunnel: w1683 -> [w2219 _]
          tunnel: w1634 -> [w2213 _]
          frame True {
            n1016 = feedback #15() -> (w2216:dbl[])  [unwired: 1 in]
            n1017 = Select(t=dbl[] [], s="R差分Bb", f=w2216) -> (s? t:f=w2215:dbl[])
            n1018 = Build Array (concatenate)(w2215, w2219) -> (w2220:dbl[])
            n1019 = feedback-in #15(w2220) -> ()
            n1020 = Index Array(array=w2220, index=w2213) -> (element=w2221:dbl)
            n1021 = Subtract(x=w2220, y=w2221) -> (x-y=→"F差分Bb":dbl[])
            n1022 = case shown="True" "R差分Bb" {
              selector: "R差分Bb" -> [_ w2223]
              frame False {
              }
              frame True {
                n1023 = Not(x=w2223) -> (.not. x?=w2222:bool)
                n1024 = local write "R差分Bb"(w2222) -> ()
              }
            }
            "N差分Bb" <- w2219
          }
          frame False {
          }
        }
        n1025 = case shown="True" w1711 {
          tunnel: w1692 -> [w2238 _]
          tunnel: w1634 -> [w2232 _]
          frame True {
            n1026 = feedback #16() -> (w2236:dbl[])  [unwired: 1 in]
            n1027 = Select(t=dbl[] [], s="R差分Cb", f=w2236) -> (s? t:f=w2235:dbl[])
            n1028 = Build Array (concatenate)(w2235, w2238) -> (w2239:dbl[])
            n1029 = feedback-in #16(w2239) -> ()
            n1030 = Index Array(array=w2239, index=w2232) -> (element=w2240:dbl)
            n1031 = Subtract(x=w2239, y=w2240) -> (x-y=→"F差分Cb":dbl[])
            n1032 = case shown="True" "R差分Cb" {
              selector: "R差分Cb" -> [_ w2242]
              frame False {
              }
              frame True {
                n1033 = Not(x=w2242) -> (.not. x?=w2241:bool)
                n1034 = local write "R差分Cb"(w2241) -> ()
              }
            }
            "N差分Cb" <- w2238
          }
          frame False {
          }
        }
        n1035 = case shown="True" w1700 {
          tunnel: w1647 -> [w2278 _]
          tunnel: w1644 -> [w2275 _]
          tunnel: w1634 -> [w2273 _]
          frame True {
            n1036 = Build Array(w2278) -> (w2274:dbl[])
            n1037 = call "绘图-分段颜色-差分.vi"("分段颜色"=w2275, "基准索引"=w2273, "光谱值"=w2274, "清空"="R差分Aa") -> ("数组"=→"F差分Aa":dbl[][])  [unwired: 7 in]
            n1038 = case shown="True" "R差分Aa" {
              selector: "R差分Aa" -> [_ w2280]
              frame False {
              }
              frame True {
                n1039 = Not(x=w2280) -> (.not. x?=w2279:bool)
                n1040 = local write "R差分Aa"(w2279) -> ()
              }
            }
            "N差分Aa" <- w2278
          }
          frame False {
          }
        }
        n1041 = call <vilib>:"Add State(s) to Queue__JKI_lib_State_Machine.vi"("State(s) in (\"\")"=w1720) -> ("States Out"=w1721:string)  [unwired: 14 in]
      }
      frame "UI: Update Graph_Diff_LT2" {
        # "长期-差分1"
        n1042 = Unbundle By Name(w2365) -> ("Time and Data.当前运行信息.当前索引子集"=w2283:i8[], "Indicators.图表相关.分段颜色"=w2284:enum32{"蓝色", "红色"}, "Time and Data.Data"=w2366:dbl[], "Sample Settings.校准.温度校准值"=w2292:dbl[], "Indicators.图表相关.基准索引"=w2281:i32)
        n1043 = Index Array(array=w2283) -> (element=w2282:i8)  [unwired: 1 in]
        n1044 = Index Array(array=w2366) -> (element #1=w2291:dbl, element #2=w2290:dbl, element #3=w2289:dbl, element #4=w2288:dbl, element #5=w2287:dbl, element #6=w2286:dbl, element #7=w2285:dbl)  [unwired: 7 in]
        n1045 = case shown="20" "差分Db" {
          tunnel: w2291 -> [w2665 w2667 w2669 w2671 _ _ _ _ _ _ w2685 w2687 _ _ _ _ _ _ _ _ _]
          tunnel: w2290 -> [w2664 _ _ _ w2673 w2675 w2677 _ _ _ _ _ w2689 w2691 _ _ _ _ _ _ _]
          tunnel: w2289 -> [_ w2666 _ _ w2672 _ _ w2679 w2681 _ _ _ _ _ w2693 w2695 _ _ _ _ _]
          tunnel: w2288 -> [_ _ w2668 _ _ w2674 _ w2678 _ w2683 _ _ _ _ _ _ w2697 w2699 _ _ _]
          tunnel: [w2665 w2667 w2669 w2671 w2673 w2675 w2677 w2679 w2681 w2683 w2685 w2687 w2689 w2691 w2693 w2695 w2697 w2699 w2701 w2703 w2705] -> w2316
          tunnel: [w2664 w2666 w2668 w2670 w2672 w2674 w2676 w2678 w2680 w2682 w2684 w2686 w2688 w2690 w2692 w2694 w2696 w2698 w2700 w2702 w2704] -> w2315
          tunnel: w2287 -> [_ _ _ w2670 _ _ w2676 _ w2680 w2682 _ _ _ _ _ _ _ _ w2701 w2703 _]
          tunnel: w2286 -> [_ _ _ _ _ _ _ _ _ _ w2684 _ w2688 _ w2692 _ w2696 _ w2700 _ w2705]
          tunnel: w2285 -> [_ _ _ _ _ _ _ _ _ _ _ w2686 _ w2690 _ w2694 _ w2698 _ w2702 w2704]
          frame 0, Default {
          }
          frame 1 {
          }
          frame 2 {
          }
          frame 3 {
          }
          frame 4 {
          }
          frame 5 {
          }
          frame 6 {
          }
          frame 7 {
          }
          frame 8 {
          }
          frame 9 {
          }
          frame 10 {
          }
          frame 11 {
          }
          frame 12 {
          }
          frame 13 {
          }
          frame 14 {
          }
          frame 15 {
          }
          frame 16 {
          }
          frame 17 {
          }
          frame 18 {
          }
          frame 19 {
          }
          frame 20 {
          }
        }
        n1046 = case shown="20" "差分Ea" {
          tunnel: w2291 -> [w2581 w2583 w2585 w2587 _ _ _ _ _ _ w2601 w2603 _ _ _ _ _ _ _ _ _]
          tunnel: w2290 -> [w2580 _ _ _ w2589 w2591 w2593 _ _ _ _ _ w2605 w2607 _ _ _ _ _ _ _]
          tunnel: w2289 -> [_ w2582 _ _ w2588 _ _ w2595 w2597 _ _ _ _ _ w2609 w2611 _ _ _ _ _]
          tunnel: w2288 -> [_ _ w2584 _ _ w2590 _ w2594 _ w2599 _ _ _ _ _ _ w2613 w2615 _ _ _]
          tunnel: [w2581 w2583 w2585 w2587 w2589 w2591 w2593 w2595 w2597 w2599 w2601 w2603 w2605 w2607 w2609 w2611 w2613 w2615 w2617 w2619 w2621] -> w2311
          tunnel: [w2580 w2582 w2584 w2586 w2588 w2590 w2592 w2594 w2596 w2598 w2600 w2602 w2604 w2606 w2608 w2610 w2612 w2614 w2616 w2618 w2620] -> w2310
          tunnel: w2287 -> [_ _ _ w2586 _ _ w2592 _ w2596 w2598 _ _ _ _ _ _ _ _ w2617 w2619 _]
          tunnel: w2286 -> [_ _ _ _ _ _ _ _ _ _ w2600 _ w2604 _ w2608 _ w2612 _ w2616 _ w2621]
          tunnel: w2285 -> [_ _ _ _ _ _ _ _ _ _ _ w2602 _ w2606 _ w2610 _ w2614 _ w2618 w2620]
          frame 0, Default {
          }
          frame 1 {
          }
          frame 2 {
          }
          frame 3 {
          }
          frame 4 {
          }
          frame 5 {
          }
          frame 6 {
          }
          frame 7 {
          }
          frame 8 {
          }
          frame 9 {
          }
          frame 10 {
          }
          frame 11 {
          }
          frame 12 {
          }
          frame 13 {
          }
          frame 14 {
          }
          frame 15 {
          }
          frame 16 {
          }
          frame 17 {
          }
          frame 18 {
          }
          frame 19 {
          }
          frame 20 {
          }
        }
        n1047 = case shown="20" "差分Da" {
          tunnel: w2291 -> [w2707 w2709 w2711 w2713 _ _ _ _ _ _ w2727 w2729 _ _ _ _ _ _ _ _ _]
          tunnel: w2290 -> [w2706 _ _ _ w2715 w2717 w2719 _ _ _ _ _ w2731 w2733 _ _ _ _ _ _ _]
          tunnel: w2289 -> [_ w2708 _ _ w2714 _ _ w2721 w2723 _ _ _ _ _ w2735 w2737 _ _ _ _ _]
          tunnel: w2288 -> [_ _ w2710 _ _ w2716 _ w2720 _ w2725 _ _ _ _ _ _ w2739 w2741 _ _ _]
          tunnel: [w2707 w2709 w2711 w2713 w2715 w2717 w2719 w2721 w2723 w2725 w2727 w2729 w2731 w2733 w2735 w2737 w2739 w2741 w2743 w2745 w2747] -> w2318
          tunnel: [w2706 w2708 w2710 w2712 w2714 w2716 w2718 w2720 w2722 w2724 w2726 w2728 w2730 w2732 w2734 w2736 w2738 w2740 w2742 w2744 w2746] -> w2317
          tunnel: w2287 -> [_ _ _ w2712 _ _ w2718 _ w2722 w2724 _ _ _ _ _ _ _ _ w2743 w2745 _]
          tunnel: w2286 -> [_ _ _ _ _ _ _ _ _ _ w2726 _ w2730 _ w2734 _ w2738 _ w2742 _ w2747]
          tunnel: w2285 -> [_ _ _ _ _ _ _ _ _ _ _ w2728 _ w2732 _ w2736 _ w2740 _ w2744 w2746]
          frame 0, Default {
          }
          frame 1 {
          }
          frame 2 {
          }
          frame 3 {
          }
          frame 4 {
          }
          frame 5 {
          }
          frame 6 {
          }
          frame 7 {
          }
          frame 8 {
          }
          frame 9 {
          }
          frame 10 {
          }
          frame 11 {
          }
          frame 12 {
          }
          frame 13 {
          }
          frame 14 {
          }
          frame 15 {
          }
          frame 16 {
          }
          frame 17 {
          }
          frame 18 {
          }
          frame 19 {
          }
          frame 20 {
          }
        }
        n1048 = case shown="20" "差分Dc" {
          tunnel: w2291 -> [w2623 w2625 w2627 w2629 _ _ _ _ _ _ w2643 w2645 _ _ _ _ _ _ _ _ _]
          tunnel: w2290 -> [w2622 _ _ _ w2631 w2633 w2635 _ _ _ _ _ w2647 w2649 _ _ _ _ _ _ _]
          tunnel: w2289 -> [_ w2624 _ _ w2630 _ _ w2637 w2639 _ _ _ _ _ w2651 w2653 _ _ _ _ _]
          tunnel: w2288 -> [_ _ w2626 _ _ w2632 _ w2636 _ w2641 _ _ _ _ _ _ w2655 w2657 _ _ _]
          tunnel: [w2623 w2625 w2627 w2629 w2631 w2633 w2635 w2637 w2639 w2641 w2643 w2645 w2647 w2649 w2651 w2653 w2655 w2657 w2659 w2661 w2663] -> w2313
          tunnel: [w2622 w2624 w2626 w2628 w2630 w2632 w2634 w2636 w2638 w2640 w2642 w2644 w2646 w2648 w2650 w2652 w2654 w2656 w2658 w2660 w2662] -> w2312
          tunnel: w2287 -> [_ _ _ w2628 _ _ w2634 _ w2638 w2640 _ _ _ _ _ _ _ _ w2659 w2661 _]
          tunnel: w2286 -> [_ _ _ _ _ _ _ _ _ _ w2642 _ w2646 _ w2650 _ w2654 _ w2658 _ w2663]
          tunnel: w2285 -> [_ _ _ _ _ _ _ _ _ _ _ w2644 _ w2648 _ w2652 _ w2656 _ w2660 w2662]
          frame 0, Default {
          }
          frame 1 {
          }
          frame 2 {
          }
          frame 3 {
          }
          frame 4 {
          }
          frame 5 {
          }
          frame 6 {
          }
          frame 7 {
          }
          frame 8 {
          }
          frame 9 {
          }
          frame 10 {
          }
          frame 11 {
          }
          frame 12 {
          }
          frame 13 {
          }
          frame 14 {
          }
          frame 15 {
          }
          frame 16 {
          }
          frame 17 {
          }
          frame 18 {
          }
          frame 19 {
          }
          frame 20 {
          }
        }
        n1049 = case shown="20" "差分Fc" {
          tunnel: w2291 -> [w2371 w2373 w2375 w2377 _ _ _ _ _ _ w2391 w2393 _ _ _ _ _ _ _ _ _]
          tunnel: w2290 -> [w2370 _ _ _ w2379 w2381 w2383 _ _ _ _ _ w2395 w2397 _ _ _ _ _ _ _]
          tunnel: w2289 -> [_ w2372 _ _ w2378 _ _ w2385 w2387 _ _ _ _ _ w2399 w2401 _ _ _ _ _]
          tunnel: w2288 -> [_ _ w2374 _ _ w2380 _ w2384 _ w2389 _ _ _ _ _ _ w2403 w2405 _ _ _]
          tunnel: [w2371 w2373 w2375 w2377 w2379 w2381 w2383 w2385 w2387 w2389 w2391 w2393 w2395 w2397 w2399 w2401 w2403 w2405 w2407 w2409 w2411] -> w2297
          tunnel: [w2370 w2372 w2374 w2376 w2378 w2380 w2382 w2384 w2386 w2388 w2390 w2392 w2394 w2396 w2398 w2400 w2402 w2404 w2406 w2408 w2410] -> w2296
          tunnel: w2287 -> [_ _ _ w2376 _ _ w2382 _ w2386 w2388 _ _ _ _ _ _ _ _ w2407 w2409 _]
          tunnel: w2286 -> [_ _ _ _ _ _ _ _ _ _ w2390 _ w2394 _ w2398 _ w2402 _ w2406 _ w2411]
          tunnel: w2285 -> [_ _ _ _ _ _ _ _ _ _ _ w2392 _ w2396 _ w2400 _ w2404 _ w2408 w2410]
          frame 0, Default {
          }
          frame 1 {
          }
          frame 2 {
          }
          frame 3 {
          }
          frame 4 {
          }
          frame 5 {
          }
          frame 6 {
          }
          frame 7 {
          }
          frame 8 {
          }
          frame 9 {
          }
          frame 10 {
          }
          frame 11 {
          }
          frame 12 {
          }
          frame 13 {
          }
          frame 14 {
          }
          frame 15 {
          }
          frame 16 {
          }
          frame 17 {
          }
          frame 18 {
          }
          frame 19 {
          }
          frame 20 {
          }
        }
        n1050 = case shown="20" "差分Fb" {
          tunnel: w2291 -> [w2413 w2415 w2417 w2419 _ _ _ _ _ _ w2433 w2435 _ _ _ _ _ _ _ _ _]
          tunnel: w2290 -> [w2412 _ _ _ w2421 w2423 w2425 _ _ _ _ _ w2437 w2439 _ _ _ _ _ _ _]
          tunnel: w2289 -> [_ w2414 _ _ w2420 _ _ w2427 w2429 _ _ _ _ _ w2441 w2443 _ _ _ _ _]
          tunnel: w2288 -> [_ _ w2416 _ _ w2422 _ w2426 _ w2431 _ _ _ _ _ _ w2445 w2447 _ _ _]
          tunnel: [w2413 w2415 w2417 w2419 w2421 w2423 w2425 w2427 w2429 w2431 w2433 w2435 w2437 w2439 w2441 w2443 w2445 w2447 w2449 w2451 w2453] -> w2300
          tunnel: [w2412 w2414 w2416 w2418 w2420 w2422 w2424 w2426 w2428 w2430 w2432 w2434 w2436 w2438 w2440 w2442 w2444 w2446 w2448 w2450 w2452] -> w2299
          tunnel: w2287 -> [_ _ _ w2418 _ _ w2424 _ w2428 w2430 _ _ _ _ _ _ _ _ w2449 w2451 _]
          tunnel: w2286 -> [_ _ _ _ _ _ _ _ _ _ w2432 _ w2436 _ w2440 _ w2444 _ w2448 _ w2453]
          tunnel: w2285 -> [_ _ _ _ _ _ _ _ _ _ _ w2434 _ w2438 _ w2442 _ w2446 _ w2450 w2452]
          frame 0, Default {
          }
          frame 1 {
          }
          frame 2 {
          }
          frame 3 {
          }
          frame 4 {
          }
          frame 5 {
          }
          frame 6 {
          }
          frame 7 {
          }
          frame 8 {
          }
          frame 9 {
          }
          frame 10 {
          }
          frame 11 {
          }
          frame 12 {
          }
          frame 13 {
          }
          frame 14 {
          }
          frame 15 {
          }
          frame 16 {
          }
          frame 17 {
          }
          frame 18 {
          }
          frame 19 {
          }
          frame 20 {
          }
        }
        n1051 = case shown="20" "差分Eb" {
          tunnel: w2291 -> [w2539 w2541 w2543 w2545 _ _ _ _ _ _ w2559 w2561 _ _ _ _ _ _ _ _ _]
          tunnel: w2290 -> [w2538 _ _ _ w2547 w2549 w2551 _ _ _ _ _ w2563 w2565 _ _ _ _ _ _ _]
          tunnel: w2289 -> [_ w2540 _ _ w2546 _ _ w2553 w2555 _ _ _ _ _ w2567 w2569 _ _ _ _ _]
          tunnel: w2288 -> [_ _ w2542 _ _ w2548 _ w2552 _ w2557 _ _ _ _ _ _ w2571 w2573 _ _ _]
          tunnel: [w2539 w2541 w2543 w2545 w2547 w2549 w2551 w2553 w2555 w2557 w2559 w2561 w2563 w2565 w2567 w2569 w2571 w2573 w2575 w2577 w2579] -> w2307
          tunnel: [w2538 w2540 w2542 w2544 w2546 w2548 w2550 w2552 w2554 w2556 w2558 w2560 w2562 w2564 w2566 w2568 w2570 w2572 w2574 w2576 w2578] -> w2306
          tunnel: w2287 -> [_ _ _ w2544 _ _ w2550 _ w2554 w2556 _ _ _ _ _ _ _ _ w2575 w2577 _]
          tunnel: w2286 -> [_ _ _ _ _ _ _ _ _ _ w2558 _ w2562 _ w2566 _ w2570 _ w2574 _ w2579]
          tunnel: w2285 -> [_ _ _ _ _ _ _ _ _ _ _ w2560 _ w2564 _ w2568 _ w2572 _ w2576 w2578]
          frame 0, Default {
          }
          frame 1 {
          }
          frame 2 {
          }
          frame 3 {
          }
          frame 4 {
          }
          frame 5 {
          }
          frame 6 {
          }
          frame 7 {
          }
          frame 8 {
          }
          frame 9 {
          }
          frame 10 {
          }
          frame 11 {
          }
          frame 12 {
          }
          frame 13 {
          }
          frame 14 {
          }
          frame 15 {
          }
          frame 16 {
          }
          frame 17 {
          }
          frame 18 {
          }
          frame 19 {
          }
          frame 20 {
          }
        }
        n1052 = case shown="20" "差分Fa" {
          tunnel: w2291 -> [w2455 w2457 w2459 w2461 _ _ _ _ _ _ w2475 w2477 _ _ _ _ _ _ _ _ _]
          tunnel: w2290 -> [w2454 _ _ _ w2463 w2465 w2467 _ _ _ _ _ w2479 w2481 _ _ _ _ _ _ _]
          tunnel: w2289 -> [_ w2456 _ _ w2462 _ _ w2469 w2471 _ _ _ _ _ w2483 w2485 _ _ _ _ _]
          tunnel: w2288 -> [_ _ w2458 _ _ w2464 _ w2468 _ w2473 _ _ _ _ _ _ w2487 w2489 _ _ _]
          tunnel: [w2455 w2457 w2459 w2461 w2463 w2465 w2467 w2469 w2471 w2473 w2475 w2477 w2479 w2481 w2483 w2485 w2487 w2489 w2491 w2493 w2495] -> w2303
          tunnel: [w2454 w2456 w2458 w2460 w2462 w2464 w2466 w2468 w2470 w2472 w2474 w2476 w2478 w2480 w2482 w2484 w2486 w2488 w2490 w2492 w2494] -> w2302
          tunnel: w2287 -> [_ _ _ w2460 _ _ w2466 _ w2470 w2472 _ _ _ _ _ _ _ _ w2491 w2493 _]
          tunnel: w2286 -> [_ _ _ _ _ _ _ _ _ _ w2474 _ w2478 _ w2482 _ w2486 _ w2490 _ w2495]
          tunnel: w2285 -> [_ _ _ _ _ _ _ _ _ _ _ w2476 _ w2480 _ w2484 _ w2488 _ w2492 w2494]
          frame 0, Default {
          }
          frame 1 {
          }
          frame 2 {
          }
          frame 3 {
          }
          frame 4 {
          }
          frame 5 {
          }
          frame 6 {
          }
          frame 7 {
          }
          frame 8 {
          }
          frame 9 {
          }
          frame 10 {
          }
          frame 11 {
          }
          frame 12 {
          }
          frame 13 {
          }
          frame 14 {
          }
          frame 15 {
          }
          frame 16 {
          }
          frame 17 {
          }
          frame 18 {
          }
          frame 19 {
          }
          frame 20 {
          }
        }
        n1053 = case shown="20" "差分Ec" {
          tunnel: w2291 -> [w2497 w2499 w2501 w2503 _ _ _ _ _ _ w2517 w2519 _ _ _ _ _ _ _ _ _]
          tunnel: w2290 -> [w2496 _ _ _ w2505 w2507 w2509 _ _ _ _ _ w2521 w2523 _ _ _ _ _ _ _]
          tunnel: w2289 -> [_ w2498 _ _ w2504 _ _ w2511 w2513 _ _ _ _ _ w2525 w2527 _ _ _ _ _]
          tunnel: w2288 -> [_ _ w2500 _ _ w2506 _ w2510 _ w2515 _ _ _ _ _ _ w2529 w2531 _ _ _]
          tunnel: [w2497 w2499 w2501 w2503 w2505 w2507 w2509 w2511 w2513 w2515 w2517 w2519 w2521 w2523 w2525 w2527 w2529 w2531 w2533 w2535 w2537] -> w2305
          tunnel: [w2496 w2498 w2500 w2502 w2504 w2506 w2508 w2510 w2512 w2514 w2516 w2518 w2520 w2522 w2524 w2526 w2528 w2530 w2532 w2534 w2536] -> w2304
          tunnel: w2287 -> [_ _ _ w2502 _ _ w2508 _ w2512 w2514 _ _ _ _ _ _ _ _ w2533 w2535 _]
          tunnel: w2286 -> [_ _ _ _ _ _ _ _ _ _ w2516 _ w2520 _ w2524 _ w2528 _ w2532 _ w2537]
          tunnel: w2285 -> [_ _ _ _ _ _ _ _ _ _ _ w2518 _ w2522 _ w2526 _ w2530 _ w2534 w2536]
          frame 0, Default {
          }
          frame 1 {
          }
          frame 2 {
          }
          frame 3 {
          }
          frame 4 {
          }
          frame 5 {
          }
          frame 6 {
          }
          frame 7 {
          }
          frame 8 {
          }
          frame 9 {
          }
          frame 10 {
          }
          frame 11 {
          }
          frame 12 {
          }
          frame 13 {
          }
          frame 14 {
          }
          frame 15 {
          }
          frame 16 {
          }
          frame 17 {
          }
          frame 18 {
          }
          frame 19 {
          }
          frame 20 {
          }
        }
        n1054 = xnode "公式 Db"("X1"=w2316, "X2"=w2315) -> ("结果"=w2325:dbl)  [unwired: 1 in, 1 out]
        n1055 = xnode "公式 Dc"("X1"=w2313, "X2"=w2312) -> ("结果"=w2328:dbl)  [unwired: 1 in, 1 out]
        n1056 = xnode "公式 Ea"("X1"=w2311, "X2"=w2310) -> ("结果"=w2331:dbl)  [unwired: 1 in, 1 out]
        n1057 = xnode "公式 Eb"("X1"=w2307, "X2"=w2306) -> ("结果"=w2334:dbl)  [unwired: 1 in, 1 out]
        n1058 = xnode "公式 Ec"("X1"=w2305, "X2"=w2304) -> ("结果"=w2337:dbl)  [unwired: 1 in, 1 out]
        n1059 = xnode "公式 Fa"("X1"=w2303, "X2"=w2302) -> ("结果"=w2340:dbl)  [unwired: 1 in, 1 out]
        n1060 = xnode "公式 Fb"("X1"=w2300, "X2"=w2299) -> ("结果"=w2343:dbl)  [unwired: 1 in, 1 out]
        n1061 = xnode "公式 Fc"("X1"=w2297, "X2"=w2296) -> ("结果"=w2346:dbl)  [unwired: 1 in, 1 out]
        n1062 = xnode "公式 Da"("X1"=w2318, "X2"=w2317) -> ("结果"=w2322:dbl)  [unwired: 1 in, 1 out]
        n1063 = Index Array(array=w2292, index="差分Db") -> (element=w2324:dbl)
        n1064 = Index Array(array=w2292, index="差分Da") -> (element=w2321:dbl)
        n1065 = Index Array(array=w2292, index="差分Dc") -> (element=w2327:dbl)
        n1066 = Index Array(array=w2292, index="差分Ea") -> (element=w2330:dbl)
        n1067 = Index Array(array=w2292, index="差分Eb") -> (element=w2333:dbl)
        n1068 = Index Array(array=w2292, index="差分Ec") -> (element=w2336:dbl)
        n1069 = Index Array(array=w2292, index="差分Fa") -> (element=w2339:dbl)
        n1070 = Index Array(array=w2292, index="差分Fb") -> (element=w2342:dbl)
        n1071 = Index Array(array=w2292, index="差分Fc") -> (element=w2345:dbl)
        n1072 = Subtract(x=w2340, y=w2339) -> (x-y=w2338:dbl)
        n1073 = Subtract(x=w2325, y=w2324) -> (x-y=w2323:dbl)
        n1074 = Subtract(x=w2334, y=w2333) -> (x-y=w2332:dbl)
        n1075 = Subtract(x=w2322, y=w2321) -> (x-y=w2320:dbl)
        n1076 = Subtract(x=w2328, y=w2327) -> (x-y=w2326:dbl)
        n1077 = Subtract(x=w2346, y=w2345) -> (x-y=w2344:dbl)
        n1078 = Subtract(x=w2331, y=w2330) -> (x-y=w2329:dbl)
        n1079 = Subtract(x=w2337, y=w2336) -> (x-y=w2335:dbl)
        n1080 = Subtract(x=w2343, y=w2342) -> (x-y=w2341:dbl)
        n1081 = Equal?(x=w2282, y="W差分Db") -> (x = y?=w2362:bool)
        n1082 = Equal?(x=w2282, y="W差分Da") -> (x = y?=w2364:bool)
        n1083 = Equal?(x=w2282, y="W差分Dc") -> (x = y?=w2361:bool)
        n1084 = Equal?(x=w2282, y="W差分Ea") -> (x = y?=w2358:bool)
        n1085 = Equal?(x=w2282, y="W差分Eb") -> (x = y?=w2357:bool)
        n1086 = Equal?(x=w2282, y="W差分Ec") -> (x = y?=w2356:bool)
        n1087 = Equal?(x=w2282, y="W差分Fa") -> (x = y?=w2355:bool)
        n1088 = Equal?(x=w2282, y="W差分Fb") -> (x = y?=w2352:bool)
        n1089 = Equal?(x=w2282, y="W差分Fc") -> (x = y?=w2350:bool)
        n1090 = case shown="True" w2362 {
          tunnel: w2323 -> [w2915 _]
          tunnel: w2281 -> [w2909 _]
          frame True {
            n1091 = feedback #17() -> (w2912:dbl[])  [unwired: 1 in]
            n1092 = Select(t=dbl[] [], s="R差分Db", f=w2912) -> (s? t:f=w2911:dbl[])
            n1093 = Build Array (concatenate)(w2911, w2915) -> (w2916:dbl[])
            n1094 = feedback-in #17(w2916) -> ()
            n1095 = Index Array(array=w2916, index=w2909) -> (element=w2917:dbl)
            n1096 = Subtract(x=w2916, y=w2917) -> (x-y=→"F差分Db":dbl[])
            n1097 = case shown="True" "R差分Db" {
              selector: "R差分Db" -> [_ w2919]
              frame False {
              }
              frame True {
                n1098 = Not(x=w2919) -> (.not. x?=w2918:bool)
                n1099 = local write "R差分Db"(w2918) -> ()
              }
            }
            "N差分Db" <- w2915
          }
          frame False {
          }
        }
        n1100 = case shown="True" w2364 {
          tunnel: w2320 -> [w2924 _]
          tunnel: w2284 -> [w2923 _]
          tunnel: w2281 -> [w2920 _]
          frame True {
            n1101 = Build Array(w2924) -> (w2921:dbl[])
            n1102 = call "绘图-分段颜色-差分.vi"("分段颜色"=w2923, "基准索引"=w2920, "光谱值"=w2921, "清空"="R差分Da") -> ("数组"=→"F差分Da":dbl[][])  [unwired: 7 in]
            n1103 = case shown="True" "R差分Da" {
              selector: "R差分Da" -> [_ w2927]
              frame False {
              }
              frame True {
                n1104 = Not(x=w2927) -> (.not. x?=w2926:bool)
                n1105 = local write "R差分Da"(w2926) -> ()
              }
            }
            "N差分Da" <- w2924
          }
          frame False {
          }
        }
        n1106 = case shown="True" w2361 {
          tunnel: w2326 -> [w2904 _]
          tunnel: w2281 -> [w2898 _]
          frame True {
            n1107 = feedback #18() -> (w2901:dbl[])  [unwired: 1 in]
            n1108 = Select(t=dbl[] [], s="R差分Dc", f=w2901) -> (s? t:f=w2900:dbl[])
            n1109 = Build Array (concatenate)(w2900, w2904) -> (w2905:dbl[])
            n1110 = feedback-in #18(w2905) -> ()
            n1111 = Index Array(array=w2905, index=w2898) -> (element=w2906:dbl)
            n1112 = Subtract(x=w2905, y=w2906) -> (x-y=→"F差分Dc":dbl[])
            n1113 = case shown="True" "R差分Dc" {
              selector: "R差分Dc" -> [_ w2908]
              frame False {
              }
              frame True {
                n1114 = Not(x=w2908) -> (.not. x?=w2907:bool)
                n1115 = local write "R差分Dc"(w2907) -> ()
              }
            }
            "N差分Dc" <- w2904
          }
          frame False {
          }
        }
        n1116 = case shown="True" w2358 {
          tunnel: w2329 -> [w2864 _]
          tunnel: w2284 -> [w2862 _]
          tunnel: w2281 -> [w2860 _]
          frame True {
            n1117 = Build Array(w2864) -> (w2861:dbl[])
            n1118 = call "绘图-分段颜色-差分.vi"("分段颜色"=w2862, "基准索引"=w2860, "光谱值"=w2861, "清空"="R差分Ea") -> ("数组"=→"F差分Ea":dbl[][])  [unwired: 7 in]
            n1119 = case shown="True" "R差分Ea" {
              selector: "R差分Ea" -> [_ w2867]
              frame False {
              }
              frame True {
                n1120 = Not(x=w2867) -> (.not. x?=w2866:bool)
                n1121 = local write "R差分Ea"(w2866) -> ()
              }
            }
            "N差分Ea" <- w2864
          }
          frame False {
          }
        }
        n1122 = case shown="True" w2357 {
          tunnel: w2332 -> [w2845 _]
          tunnel: w2281 -> [w2839 _]
          frame True {
            n1123 = feedback #19() -> (w2842:dbl[])  [unwired: 1 in]
            n1124 = Select(t=dbl[] [], s="R差分Eb", f=w2842) -> (s? t:f=w2841:dbl[])
            n1125 = Build Array (concatenate)(w2841, w2845) -> (w2846:dbl[])
            n1126 = feedback-in #19(w2846) -> ()
            n1127 = Index Array(array=w2846, index=w2839) -> (element=w2847:dbl)
            n1128 = Subtract(x=w2846, y=w2847) -> (x-y=→"F差分Eb":dbl[])
            n1129 = case shown="True" "R差分Eb" {
              selector: "R差分Eb" -> [_ w2849]
              frame False {
              }
              frame True {
                n1130 = Not(x=w2849) -> (.not. x?=w2848:bool)
                n1131 = local write "R差分Eb"(w2848) -> ()
              }
            }
            "N差分Eb" <- w2845
          }
          frame False {
          }
        }
        n1132 = case shown="True" w2356 {
          tunnel: w2335 -> [w2824 _]
          tunnel: w2281 -> [w2818 _]
          frame True {
            n1133 = feedback #20() -> (w2821:dbl[])  [unwired: 1 in]
            n1134 = Select(t=dbl[] [], s="R差分Ec", f=w2821) -> (s? t:f=w2820:dbl[])
            n1135 = Build Array (concatenate)(w2820, w2824) -> (w2825:dbl[])
            n1136 = feedback-in #20(w2825) -> ()
            n1137 = Index Array(array=w2825, index=w2818) -> (element=w2826:dbl)
            n1138 = Subtract(x=w2825, y=w2826) -> (x-y=→"F差分Ec":dbl[])
            n1139 = case shown="True" "R差分Ec" {
              selector: "R差分Ec" -> [_ w2828]
              frame False {
              }
              frame True {
                n1140 = Not(x=w2828) -> (.not. x?=w2827:bool)
                n1141 = local write "R差分Ec"(w2827) -> ()
              }
            }
            "N差分Ec" <- w2824
          }
          frame False {
          }
        }
        n1142 = case shown="True" w2355 {
          tunnel: w2338 -> [w2803 _]
          tunnel: w2284 -> [w2802 _]
          tunnel: w2281 -> [w2800 _]
          frame True {
            n1143 = Build Array(w2803) -> (w2801:dbl[])
            n1144 = call "绘图-分段颜色-差分.vi"("分段颜色"=w2802, "基准索引"=w2800, "光谱值"=w2801, "清空"="R差分Fa") -> ("数组"=→"F差分Fa":dbl[][])  [unwired: 7 in]
            n1145 = case shown="True" "R差分Fa" {
              selector: "R差分Fa" -> [_ w2807]
              frame False {
              }
              frame True {
                n1146 = Not(x=w2807) -> (.not. x?=w2806:bool)
                n1147 = local write "R差分Fa"(w2806) -> ()
              }
            }
            "N差分Fa" <- w2803
          }
          frame False {
          }
        }
        n1148 = case shown="True" w2352 {
          tunnel: w2341 -> [w2785 _]
          tunnel: w2281 -> [w2779 _]
          frame True {
            n1149 = feedback #21() -> (w2782:dbl[])  [unwired: 1 in]
            n1150 = Select(t=dbl[] [], s="R差分Fb", f=w2782) -> (s? t:f=w2781:dbl[])
            n1151 = Build Array (concatenate)(w2781, w2785) -> (w2786:dbl[])
            n1152 = feedback-in #21(w2786) -> ()
            n1153 = Index Array(array=w2786, index=w2779) -> (element=w2787:dbl)
            n1154 = case shown="True" "R差分Fb" {
              selector: "R差分Fb" -> [_ w2789]
              frame False {
              }
              frame True {
                n1155 = Not(x=w2789) -> (.not. x?=w2788:bool)
                n1156 = local write "R差分Fb"(w2788) -> ()
              }
            }
            n1157 = Subtract(x=w2786, y=w2787) -> (x-y=→"F差分Fb":dbl[])
            "N差分Fb" <- w2785
          }
          frame False {
          }
        }
        n1158 = case shown="True" w2350 {
          tunnel: w2344 -> [w2764 _]
          tunnel: w2281 -> [w2758 _]
          frame True {
            n1159 = feedback #22() -> (w2761:dbl[])  [unwired: 1 in]
            n1160 = Select(t=dbl[] [], s="R差分Fc", f=w2761) -> (s? t:f=w2760:dbl[])
            n1161 = Build Array (concatenate)(w2760, w2764) -> (w2765:dbl[])
            n1162 = feedback-in #22(w2765) -> ()
            n1163 = Index Array(array=w2765, index=w2758) -> (element=w2766:dbl)
            n1164 = Subtract(x=w2765, y=w2766) -> (x-y=→"F差分Fc":dbl[])
            n1165 = case shown="True" "R差分Fc" {
              selector: "R差分Fc" -> [_ w2768]
              frame False {
              }
              frame True {
                n1166 = Not(x=w2768) -> (.not. x?=w2767:bool)
                n1167 = local write "R差分Fc"(w2767) -> ()
              }
            }
            "N差分Fc" <- w2764
          }
          frame False {
          }
        }
        n1168 = call <vilib>:"Add State(s) to Queue__JKI_lib_State_Machine.vi"("State(s) in (\"\")"=w2367) -> ("States Out"=w2368:string)  [unwired: 14 in]
      }
      frame "UI: Update Graph_Diff_LT3" {
        # "长期-差分1"
        n1169 = Unbundle By Name(w2940) -> ("Time and Data.当前运行信息.当前索引子集"=w2939:i8[], "Indicators.图表相关.分段颜色"=w2938:enum32{"蓝色", "红色"}, "Time and Data.Data"=w2941:dbl[], "Sample Settings.校准.温度校准值"=w2930:dbl[], "Indicators.图表相关.基准索引"=w2928:i32)
        n1170 = Index Array(array=w2939) -> (element=w2929:i8)  [unwired: 1 in]
        n1171 = Index Array(array=w2941) -> (element #1=w2937:dbl, element #2=w2936:dbl, element #3=w2935:dbl, element #4=w2934:dbl, element #5=w2933:dbl, element #6=w2932:dbl, element #7=w2931:dbl)  [unwired: 7 in]
        n1172 = case shown="20" "差分Gc" {
          tunnel: w2937 -> [w3180 w3182 w3184 w3186 _ _ _ _ _ _ w3200 w3202 _ _ _ _ _ _ _ _ _]
          tunnel: w2936 -> [w3179 _ _ _ w3188 w3190 w3192 _ _ _ _ _ w3204 w3206 _ _ _ _ _ _ _]
          tunnel: w2935 -> [_ w3181 _ _ w3187 _ _ w3194 w3196 _ _ _ _ _ w3208 w3210 _ _ _ _ _]
          tunnel: w2934 -> [_ _ w3183 _ _ w3189 _ w3193 _ w3198 _ _ _ _ _ _ w3212 w3214 _ _ _]
          tunnel: [w3180 w3182 w3184 w3186 w3188 w3190 w3192 w3194 w3196 w3198 w3200 w3202 w3204 w3206 w3208 w3210 w3212 w3214 w3216 w3218 w3220] -> w2973
          tunnel: [w3179 w3181 w3183 w3185 w3187 w3189 w3191 w3193 w3195 w3197 w3199 w3201 w3203 w3205 w3207 w3209 w3211 w3213 w3215 w3217 w3219] -> w2972
          tunnel: w2933 -> [_ _ _ w3185 _ _ w3191 _ w3195 w3197 _ _ _ _ _ _ _ _ w3216 w3218 _]
          tunnel: w2932 -> [_ _ _ _ _ _ _ _ _ _ w3199 _ w3203 _ w3207 _ w3211 _ w3215 _ w3220]
          tunnel: w2931 -> [_ _ _ _ _ _ _ _ _ _ _ w3201 _ w3205 _ w3209 _ w3213 _ w3217 w3219]
          frame 0, Default {
          }
          frame 1 {
          }
          frame 2 {
          }
          frame 3 {
          }
          frame 4 {
          }
          frame 5 {
          }
          frame 6 {
          }
          frame 7 {
          }
          frame 8 {
          }
          frame 9 {
          }
          frame 10 {
          }
          frame 11 {
          }
          frame 12 {
          }
          frame 13 {
          }
          frame 14 {
          }
          frame 15 {
          }
          frame 16 {
          }
          frame 17 {
          }
          frame 18 {
          }
          frame 19 {
          }
          frame 20 {
          }
        }
        n1173 = case shown="20" "差分Hc" {
          tunnel: w2937 -> [w2994 w2996 w2998 w3000 _ _ _ _ _ _ w3014 w3016 _ _ _ _ _ _ _ _ _]
          tunnel: w2936 -> [w2993 _ _ _ w3002 w3004 w3006 _ _ _ _ _ w3018 w3020 _ _ _ _ _ _ _]
          tunnel: w2935 -> [_ w2995 _ _ w3001 _ _ w3008 w3010 _ _ _ _ _ w3022 w3024 _ _ _ _ _]
          tunnel: w2934 -> [_ _ w2997 _ _ w3003 _ w3007 _ w3012 _ _ _ _ _ _ w3026 w3028 _ _ _]
          tunnel: [w2994 w2996 w2998 w3000 w3002 w3004 w3006 w3008 w3010 w3012 w3014 w3016 w3018 w3020 w3022 w3024 w3026 w3028 w3030 w3032 w3034] -> w2949
          tunnel: [w2993 w2995 w2997 w2999 w3001 w3003 w3005 w3007 w3009 w3011 w3013 w3015 w3017 w3019 w3021 w3023 w3025 w3027 w3029 w3031 w3033] -> w2948
          tunnel: w2933 -> [_ _ _ w2999 _ _ w3005 _ w3009 w3011 _ _ _ _ _ _ _ _ w3030 w3032 _]
          tunnel: w2932 -> [_ _ _ _ _ _ _ _ _ _ w3013 _ w3017 _ w3021 _ w3025 _ w3029 _ w3034]
          tunnel: w2931 -> [_ _ _ _ _ _ _ _ _ _ _ w3015 _ w3019 _ w3023 _ w3027 _ w3031 w3033]
          frame 0, Default {
          }
          frame 1 {
          }
          frame 2 {
          }
          frame 3 {
          }
          frame 4 {
          }
          frame 5 {
          }
          frame 6 {
          }
          frame 7 {
          }
          frame 8 {
          }
          frame 9 {
          }
          frame 10 {
          }
          frame 11 {
          }
          frame 12 {
          }
          frame 13 {
          }
          frame 14 {
          }
          frame 15 {
          }
          frame 16 {
          }
          frame 17 {
          }
          frame 18 {
          }
          frame 19 {
          }
          frame 20 {
          }
        }
        n1174 = case shown="20" "差分Gb" {
          tunnel: w2937 -> [w3222 w3224 w3226 w3228 _ _ _ _ _ _ w3242 w3244 _ _ _ _ _ _ _ _ _]
          tunnel: w2936 -> [w3221 _ _ _ w3230 w3232 w3234 _ _ _ _ _ w3246 w3248 _ _ _ _ _ _ _]
          tunnel: w2935 -> [_ w3223 _ _ w3229 _ _ w3236 w3238 _ _ _ _ _ w3250 w3252 _ _ _ _ _]
          tunnel: w2934 -> [_ _ w3225 _ _ w3231 _ w3235 _ w3240 _ _ _ _ _ _ w3254 w3256 _ _ _]
          tunnel: [w3222 w3224 w3226 w3228 w3230 w3232 w3234 w3236 w3238 w3240 w3242 w3244 w3246 w3248 w3250 w3252 w3254 w3256 w3258 w3260 w3262] -> w2975
          tunnel: [w3221 w3223 w3225 w3227 w3229 w3231 w3233 w3235 w3237 w3239 w3241 w3243 w3245 w3247 w3249 w3251 w3253 w3255 w3257 w3259 w3261] -> w2974
          tunnel: w2933 -> [_ _ _ w3227 _ _ w3233 _ w3237 w3239 _ _ _ _ _ _ _ _ w3258 w3260 _]
          tunnel: w2932 -> [_ _ _ _ _ _ _ _ _ _ w3241 _ w3245 _ w3249 _ w3253 _ w3257 _ w3262]
          tunnel: w2931 -> [_ _ _ _ _ _ _ _ _ _ _ w3243 _ w3247 _ w3251 _ w3255 _ w3259 w3261]
          frame 0, Default {
          }
          frame 1 {
          }
          frame 2 {
          }
          frame 3 {
          }
          frame 4 {
          }
          frame 5 {
          }
          frame 6 {
          }
          frame 7 {
          }
          frame 8 {
          }
          frame 9 {
          }
          frame 10 {
          }
          frame 11 {
          }
          frame 12 {
          }
          frame 13 {
          }
          frame 14 {
          }
          frame 15 {
          }
          frame 16 {
          }
          frame 17 {
          }
          frame 18 {
          }
          frame 19 {
          }
          frame 20 {
          }
        }
        n1175 = case shown="20" "差分Hb" {
          tunnel: w2937 -> [w3036 w3038 w3040 w3042 _ _ _ _ _ _ w3056 w3058 _ _ _ _ _ _ _ _ _]
          tunnel: w2936 -> [w3035 _ _ _ w3044 w3046 w3048 _ _ _ _ _ w3060 w3062 _ _ _ _ _ _ _]
          tunnel: w2935 -> [_ w3037 _ _ w3043 _ _ w3050 w3052 _ _ _ _ _ w3064 w3066 _ _ _ _ _]
          tunnel: w2934 -> [_ _ w3039 _ _ w3045 _ w3049 _ w3054 _ _ _ _ _ _ w3068 w3070 _ _ _]
          tunnel: [w3036 w3038 w3040 w3042 w3044 w3046 w3048 w3050 w3052 w3054 w3056 w3058 w3060 w3062 w3064 w3066 w3068 w3070 w3072 w3074 w3076] -> w2951
          tunnel: [w3035 w3037 w3039 w3041 w3043 w3045 w3047 w3049 w3051 w3053 w3055 w3057 w3059 w3061 w3063 w3065 w3067 w3069 w3071 w3073 w3075] -> w2950
          tunnel: w2933 -> [_ _ _ w3041 _ _ w3047 _ w3051 w3053 _ _ _ _ _ _ _ _ w3072 w3074 _]
          tunnel: w2932 -> [_ _ _ _ _ _ _ _ _ _ w3055 _ w3059 _ w3063 _ w3067 _ w3071 _ w3076]
          tunnel: w2931 -> [_ _ _ _ _ _ _ _ _ _ _ w3057 _ w3061 _ w3065 _ w3069 _ w3073 w3075]
          frame 0, Default {
          }
          frame 1 {
          }
          frame 2 {
          }
          frame 3 {
          }
          frame 4 {
          }
          frame 5 {
          }
          frame 6 {
          }
          frame 7 {
          }
          frame 8 {
          }
          frame 9 {
          }
          frame 10 {
          }
          frame 11 {
          }
          frame 12 {
          }
          frame 13 {
          }
          frame 14 {
          }
          frame 15 {
          }
          frame 16 {
          }
          frame 17 {
          }
          frame 18 {
          }
          frame 19 {
          }
          frame 20 {
          }
        }
        n1176 = case shown="20" "差分Ga" {
          tunnel: w2937 -> [w3264 w3266 w3268 w3270 _ _ _ _ _ _ w3284 w3286 _ _ _ _ _ _ _ _ _]
          tunnel: w2936 -> [w3263 _ _ _ w3272 w3274 w3276 _ _ _ _ _ w3288 w3290 _ _ _ _ _ _ _]
          tunnel: w2935 -> [_ w3265 _ _ w3271 _ _ w3278 w3280 _ _ _ _ _ w3292 w3294 _ _ _ _ _]
          tunnel: w2934 -> [_ _ w3267 _ _ w3273 _ w3277 _ w3282 _ _ _ _ _ _ w3296 w3298 _ _ _]
          tunnel: [w3264 w3266 w3268 w3270 w3272 w3274 w3276 w3278 w3280 w3282 w3284 w3286 w3288 w3290 w3292 w3294 w3296 w3298 w3300 w3302 w3304] -> w2977
          tunnel: [w3263 w3265 w3267 w3269 w3271 w3273 w3275 w3277 w3279 w3281 w3283 w3285 w3287 w3289 w3291 w3293 w3295 w3297 w3299 w3301 w3303] -> w2976
          tunnel: w2933 -> [_ _ _ w3269 _ _ w3275 _ w3279 w3281 _ _ _ _ _ _ _ _ w3300 w3302 _]
          tunnel: w2932 -> [_ _ _ _ _ _ _ _ _ _ w3283 _ w3287 _ w3291 _ w3295 _ w3299 _ w3304]
          tunnel: w2931 -> [_ _ _ _ _ _ _ _ _ _ _ w3285 _ w3289 _ w3293 _ w3297 _ w3301 w3303]
          frame 0, Default {
          }
          frame 1 {
          }
          frame 2 {
          }
          frame 3 {
          }
          frame 4 {
          }
          frame 5 {
          }
          frame 6 {
          }
          frame 7 {
          }
          frame 8 {
          }
          frame 9 {
          }
          frame 10 {
          }
          frame 11 {
          }
          frame 12 {
          }
          frame 13 {
          }
          frame 14 {
          }
          frame 15 {
          }
          frame 16 {
          }
          frame 17 {
          }
          frame 18 {
          }
          frame 19 {
          }
          frame 20 {
          }
        }
        n1177 = case shown="20" "差分Ha" {
          tunnel: w2937 -> [w3078 w3080 w3082 w3084 _ _ _ _ _ _ w3098 w3100 _ _ _ _ _ _ _ _ _]
          tunnel: w2936 -> [w3077 _ _ _ w3086 w3088 w3090 _ _ _ _ _ w3102 w3104 _ _ _ _ _ _ _]
          tunnel: w2935 -> [_ w3079 _ _ w3085 _ _ w3092 w3094 _ _ _ _ _ w3106 w3108 _ _ _ _ _]
          tunnel: w2934 -> [_ _ w3081 _ _ w3087 _ w3091 _ w3096 _ _ _ _ _ _ w3110 w3112 _ _ _]
          tunnel: [w3078 w3080 w3082 w3084 w3086 w3088 w3090 w3092 w3094 w3096 w3098 w3100 w3102 w3104 w3106 w3108 w3110 w3112 w3114 w3116 w3118] -> w2953
          tunnel: [w3077 w3079 w3081 w3083 w3085 w3087 w3089 w3091 w3093 w3095 w3097 w3099 w3101 w3103 w3105 w3107 w3109 w3111 w3113 w3115 w3117] -> w2952
          tunnel: w2933 -> [_ _ _ w3083 _ _ w3089 _ w3093 w3095 _ _ _ _ _ _ _ _ w3114 w3116 _]
          tunnel: w2932 -> [_ _ _ _ _ _ _ _ _ _ w3097 _ w3101 _ w3105 _ w3109 _ w3113 _ w3118]
          tunnel: w2931 -> [_ _ _ _ _ _ _ _ _ _ _ w3099 _ w3103 _ w3107 _ w3111 _ w3115 w3117]
          frame 0, Default {
          }
          frame 1 {
          }
          frame 2 {
          }
          frame 3 {
          }
          frame 4 {
          }
          frame 5 {
          }
          frame 6 {
          }
          frame 7 {
          }
          frame 8 {
          }
          frame 9 {
          }
          frame 10 {
          }
          frame 11 {
          }
          frame 12 {
          }
          frame 13 {
          }
          frame 14 {
          }
          frame 15 {
          }
          frame 16 {
          }
          frame 17 {
          }
          frame 18 {
          }
          frame 19 {
          }
          frame 20 {
          }
        }
        n1178 = xnode "公式 Ga"("X1"=w2977, "X2"=w2976) -> ("结果"=w2980:dbl)  [unwired: 1 in, 1 out]
        n1179 = xnode "公式 Ha"("X1"=w2953, "X2"=w2952) -> ("结果"=w2956:dbl)  [unwired: 1 in, 1 out]
        n1180 = xnode "公式 Gb"("X1"=w2975, "X2"=w2974) -> ("结果"=w2983:dbl)  [unwired: 1 in, 1 out]
        n1181 = xnode "公式 Gc"("X1"=w2973, "X2"=w2972) -> ("结果"=w2986:dbl)  [unwired: 1 in, 1 out]
        n1182 = xnode "公式 Hb"("X1"=w2951, "X2"=w2950) -> ("结果"=w2959:dbl)  [unwired: 1 in, 1 out]
        n1183 = xnode "公式 Hc"("X1"=w2949, "X2"=w2948) -> ("结果"=w2962:dbl)  [unwired: 1 in, 1 out]
        n1184 = Index Array(array=w2930, index="差分Ga") -> (element=w2979:dbl)
        n1185 = Index Array(array=w2930, index="差分Ha") -> (element=w2955:dbl)
        n1186 = Index Array(array=w2930, index="差分Gb") -> (element=w2982:dbl)
        n1187 = Index Array(array=w2930, index="差分Gc") -> (element=w2985:dbl)
        n1188 = Index Array(array=w2930, index="差分Hb") -> (element=w2958:dbl)
        n1189 = Index Array(array=w2930, index="差分Hc") -> (element=w2961:dbl)
        n1190 = Subtract(x=w2980, y=w2979) -> (x-y=w2978:dbl)
        n1191 = Subtract(x=w2956, y=w2955) -> (x-y=w2954:dbl)
        n1192 = Subtract(x=w2986, y=w2985) -> (x-y=w2984:dbl)
        n1193 = Subtract(x=w2962, y=w2961) -> (x-y=w2960:dbl)
        n1194 = Subtract(x=w2983, y=w2982) -> (x-y=w2981:dbl)
        n1195 = Subtract(x=w2959, y=w2958) -> (x-y=w2957:dbl)
        n1196 = Equal?(x=w2929, y="W差分Ga") -> (x = y?=w2989:bool)
        n1197 = Equal?(x=w2929, y="W差分Ha") -> (x = y?=w2965:bool)
        n1198 = Equal?(x=w2929, y="W差分Gb") -> (x = y?=w2988:bool)
        n1199 = Equal?(x=w2929, y="W差分Gc") -> (x = y?=w2987:bool)
        n1200 = Equal?(x=w2929, y="W差分Hb") -> (x = y?=w2964:bool)
        n1201 = Equal?(x=w2929, y="W差分Hc") -> (x = y?=w2963:bool)
        n1202 = case shown="True" w2989 {
          tunnel: w2978 -> [w3360 _]
          tunnel: w2938 -> [w3362 _]
          tunnel: w2928 -> [w3357 _]
          frame True {
            n1203 = Build Array(w3360) -> (w3358:dbl[])
            n1204 = call "绘图-分段颜色-差分.vi"("分段颜色"=w3362, "基准索引"=w3357, "光谱值"=w3358, "清空"="R差分Ga") -> ("数组"=→"F差分Ga":dbl[][])  [unwired: 7 in]
            n1205 = case shown="True" "R差分Ga" {
              selector: "R差分Ga" -> [_ w3364]
              frame False {
              }
              frame True {
                n1206 = Not(x=w3364) -> (.not. x?=w3363:bool)
                n1207 = local write "R差分Ga"(w3363) -> ()
              }
            }
            "N差分Ga" <- w3360
          }
          frame False {
          }
        }
        n1208 = case shown="True" w2965 {
          tunnel: w2954 -> [w3175 _]
          tunnel: w2938 -> [w3173 _]
          tunnel: w2928 -> [w3171 _]
          frame True {
            n1209 = Build Array(w3175) -> (w3172:dbl[])
            n1210 = call "绘图-分段颜色-差分.vi"("分段颜色"=w3173, "基准索引"=w3171, "光谱值"=w3172, "清空"="R差分Ha") -> ("数组"=→"F差分Ha":dbl[][])  [unwired: 7 in]
            n1211 = case shown="True" "R差分Ha" {
              selector: "R差分Ha" -> [_ w3178]
              frame False {
              }
              frame True {
                n1212 = Not(x=w3178) -> (.not. x?=w3177:bool)
                n1213 = local write "R差分Ha"(w3177) -> ()
              }
            }
            "N差分Ha" <- w3175
          }
          frame False {
          }
        }
        n1214 = case shown="True" w2988 {
          tunnel: w2981 -> [w3342 _]
          tunnel: w2928 -> [w3336 _]
          frame True {
            n1215 = feedback #23() -> (w3339:dbl[])  [unwired: 1 in]
            n1216 = Select(t=dbl[] [], s="R差分Gb", f=w3339) -> (s? t:f=w3338:dbl[])
            n1217 = Build Array (concatenate)(w3338, w3342) -> (w3343:dbl[])
            n1218 = feedback-in #23(w3343) -> ()
            n1219 = Index Array(array=w3343, index=w3336) -> (element=w3344:dbl)
            n1220 = Subtract(x=w3343, y=w3344) -> (x-y=→"F差分Gb":dbl[])
            n1221 = case shown="True" "R差分Gb" {
              selector: "R差分Gb" -> [_ w3346]
              frame False {
              }
              frame True {
                n1222 = Not(x=w3346) -> (.not. x?=w3345:bool)
                n1223 = local write "R差分Gb"(w3345) -> ()
              }
            }
            "N差分Gb" <- w3342
          }
          frame False {
          }
        }
        n1224 = case shown="True" w2987 {
          tunnel: w2984 -> [w3321 _]
          tunnel: w2928 -> [w3315 _]
          frame True {
            n1225 = feedback #24() -> (w3318:dbl[])  [unwired: 1 in]
            n1226 = Select(t=dbl[] [], s="R差分Gc", f=w3318) -> (s? t:f=w3317:dbl[])
            n1227 = Build Array (concatenate)(w3317, w3321) -> (w3322:dbl[])
            n1228 = feedback-in #24(w3322) -> ()
            n1229 = Index Array(array=w3322, index=w3315) -> (element=w3323:dbl)
            n1230 = Subtract(x=w3322, y=w3323) -> (x-y=→"F差分Gc":dbl[])
            n1231 = case shown="True" "R差分Gc" {
              selector: "R差分Gc" -> [_ w3325]
              frame False {
              }
              frame True {
                n1232 = Not(x=w3325) -> (.not. x?=w3324:bool)
                n1233 = local write "R差分Gc"(w3324) -> ()
              }
            }
            "N差分Gc" <- w3321
          }
          frame False {
          }
        }
        n1234 = case shown="True" w2964 {
          tunnel: w2957 -> [w3156 _]
          tunnel: w2928 -> [w3150 _]
          frame True {
            n1235 = feedback #25() -> (w3153:dbl[])  [unwired: 1 in]
            n1236 = Select(t=dbl[] [], s="R差分Hb", f=w3153) -> (s? t:f=w3152:dbl[])
            n1237 = Build Array (concatenate)(w3152, w3156) -> (w3157:dbl[])
            n1238 = feedback-in #25(w3157) -> ()
            n1239 = Index Array(array=w3157, index=w3150) -> (element=w3158:dbl)
            n1240 = Subtract(x=w3157, y=w3158) -> (x-y=→"F差分Hb":dbl[])
            n1241 = case shown="True" "R差分Hb" {
              selector: "R差分Hb" -> [_ w3160]
              frame False {
              }
              frame True {
                n1242 = Not(x=w3160) -> (.not. x?=w3159:bool)
                n1243 = local write "R差分Hb"(w3159) -> ()
              }
            }
            "N差分Hb" <- w3156
          }
          frame False {
          }
        }
        n1244 = case shown="True" w2963 {
          tunnel: w2960 -> [w3135 _]
          tunnel: w2928 -> [w3129 _]
          frame True {
            n1245 = feedback #26() -> (w3132:dbl[])  [unwired: 1 in]
            n1246 = Select(t=dbl[] [], s="R差分Hc", f=w3132) -> (s? t:f=w3131:dbl[])
            n1247 = Build Array (concatenate)(w3131, w3135) -> (w3136:dbl[])
            n1248 = feedback-in #26(w3136) -> ()
            n1249 = Index Array(array=w3136, index=w3129) -> (element=w3137:dbl)
            n1250 = Subtract(x=w3136, y=w3137) -> (x-y=→"F差分Hc":dbl[])
            n1251 = case shown="True" "R差分Hc" {
              selector: "R差分Hc" -> [_ w3139]
              frame False {
              }
              frame True {
                n1252 = Not(x=w3139) -> (.not. x?=w3138:bool)
                n1253 = local write "R差分Hc"(w3138) -> ()
              }
            }
            "N差分Hc" <- w3135
          }
          frame False {
          }
        }
        n1254 = call <vilib>:"Add State(s) to Queue__JKI_lib_State_Machine.vi"("State(s) in (\"\")"=w2990) -> ("States Out"=w2991:string)  [unwired: 14 in]
      }
      frame "UI: Update Graph_Diff_Wave" {
        w3384 = 1 ("长度")
        w3383 = 1 ("长度")
        w3382 = 1 ("长度")
        w3381 = 1 ("长度")
        w3380 = 1 ("长度")
        w3379 = 1 ("长度")
        n1255 = Unbundle By Name(w3378) -> ("Indicators.图表相关.分段颜色"=w3370:enum32{"蓝色", "红色"}, "Sample Settings.测量.每波长测量次数"=w3371:i32, "Time and Data.校准值.1环(校准值)"=w3377:dbl[][], "Time and Data.校准值.2环(校准值)"=w3376:dbl[][], "Time and Data.校准值.3环(校准值)"=w3368:dbl[][], "Time and Data.校准值.4环(校准值)"=w3375:dbl[][], "Time and Data.校准值.5环(校准值)"=w3374:dbl[][], "Time and Data.校准值.6环(校准值)"=w3373:dbl[][], "Time and Data.校准值.7环(校准值)"=w3372:dbl[][], "Indicators.图表相关.基准索引"=w3369:i32)
        n1256 = local write "程序状态"("周期结束" ("程序状态")) -> ()
        n1257 = case shown="19" "差分Y2" {
          tunnel: w3377 -> [w3654 w3656 w3658 w3660 _ _ _ _ _ _ w3674 w3676 _ _ _ _ _ _ _ _ _]
          tunnel: w3376 -> [w3653 _ _ _ w3662 w3664 w3666 _ _ _ _ _ w3678 w3680 _ _ _ _ _ _ _]
          tunnel: w3368 -> [_ w3655 _ _ w3661 _ _ w3668 w3670 _ _ _ _ _ w3682 w3684 _ _ _ _ _]
          tunnel: w3375 -> [_ _ w3657 _ _ w3663 _ w3667 _ w3672 _ _ _ _ _ _ w3686 w3688 _ _ _]
          tunnel: [w3654 w3656 w3658 w3660 w3662 w3664 w3666 w3668 w3670 w3672 w3674 w3676 w3678 w3680 w3682 w3684 w3686 w3688 w3690 w3692 w3694] -> w3443
          tunnel: [w3653 w3655 w3657 w3659 w3661 w3663 w3665 w3667 w3669 w3671 w3673 w3675 w3677 w3679 w3681 w3683 w3685 w3687 w3689 w3691 w3693] -> w3439
          tunnel: w3374 -> [_ _ _ w3659 _ _ w3665 _ w3669 w3671 _ _ _ _ _ _ _ _ w3690 w3692 _]
          tunnel: w3373 -> [_ _ _ _ _ _ _ _ _ _ w3673 _ w3677 _ w3681 _ w3685 _ w3689 _ w3694]
          tunnel: w3372 -> [_ _ _ _ _ _ _ _ _ _ _ w3675 _ w3679 _ w3683 _ w3687 _ w3691 w3693]
          frame 0, Default {
          }
          frame 1 {
          }
          frame 2 {
          }
          frame 3 {
          }
          frame 4 {
          }
          frame 5 {
          }
          frame 6 {
          }
          frame 7 {
          }
          frame 8 {
          }
          frame 9 {
          }
          frame 10 {
          }
          frame 11 {
          }
          frame 12 {
          }
          frame 13 {
          }
          frame 14 {
          }
          frame 15 {
          }
          frame 16 {
          }
          frame 17 {
          }
          frame 18 {
          }
          frame 19 {
          }
          frame 20 {
          }
        }
        n1258 = case shown="19" "差分Y3" {
          tunnel: w3377 -> [w3496 w3498 w3500 w3502 _ _ _ _ _ _ w3516 w3518 _ _ _ _ _ _ _ _ _]
          tunnel: w3376 -> [w3495 _ _ _ w3504 w3506 w3508 _ _ _ _ _ w3520 w3522 _ _ _ _ _ _ _]
          tunnel: w3368 -> [_ w3497 _ _ w3503 _ _ w3510 w3512 _ _ _ _ _ w3524 w3526 _ _ _ _ _]
          tunnel: w3375 -> [_ _ w3499 _ _ w3505 _ w3509 _ w3514 _ _ _ _ _ _ w3528 w3530 _ _ _]
          tunnel: [w3496 w3498 w3500 w3502 w3504 w3506 w3508 w3510 w3512 w3514 w3516 w3518 w3520 w3522 w3524 w3526 w3528 w3530 w3532 w3534 w3536] -> w3396
          tunnel: [w3495 w3497 w3499 w3501 w3503 w3505 w3507 w3509 w3511 w3513 w3515 w3517 w3519 w3521 w3523 w3525 w3527 w3529 w3531 w3533 w3535] -> w3400
          tunnel: w3374 -> [_ _ _ w3501 _ _ w3507 _ w3511 w3513 _ _ _ _ _ _ _ _ w3532 w3534 _]
          tunnel: w3373 -> [_ _ _ _ _ _ _ _ _ _ w3515 _ w3519 _ w3523 _ w3527 _ w3531 _ w3536]
          tunnel: w3372 -> [_ _ _ _ _ _ _ _ _ _ _ w3517 _ w3521 _ w3525 _ w3529 _ w3533 w3535]
          frame 0, Default {
          }
          frame 1 {
          }
          frame 2 {
          }
          frame 3 {
          }
          frame 4 {
          }
          frame 5 {
          }
          frame 6 {
          }
          frame 7 {
          }
          frame 8 {
          }
          frame 9 {
          }
          frame 10 {
          }
          frame 11 {
          }
          frame 12 {
          }
          frame 13 {
          }
          frame 14 {
          }
          frame 15 {
          }
          frame 16 {
          }
          frame 17 {
          }
          frame 18 {
          }
          frame 19 {
          }
          frame 20 {
          }
        }
        n1259 = case shown="19" "差分Y" {
          tunnel: w3377 -> [w3764 w3766 w3768 w3770 _ _ _ _ _ _ w3784 w3786 _ _ _ _ _ _ _ _ _]
          tunnel: w3376 -> [w3763 _ _ _ w3772 w3774 w3776 _ _ _ _ _ w3788 w3790 _ _ _ _ _ _ _]
          tunnel: w3368 -> [_ w3765 _ _ w3771 _ _ w3778 w3780 _ _ _ _ _ w3792 w3794 _ _ _ _ _]
          tunnel: w3375 -> [_ _ w3767 _ _ w3773 _ w3777 _ w3782 _ _ _ _ _ _ w3796 w3798 _ _ _]
          tunnel: [w3764 w3766 w3768 w3770 w3772 w3774 w3776 w3778 w3780 w3782 w3784 w3786 w3788 w3790 w3792 w3794 w3796 w3798 w3800 w3802 w3804] -> w3446
          tunnel: [w3763 w3765 w3767 w3769 w3771 w3773 w3775 w3777 w3779 w3781 w3783 w3785 w3787 w3789 w3791 w3793 w3795 w3797 w3799 w3801 w3803] -> w3450
          tunnel: w3374 -> [_ _ _ w3769 _ _ w3775 _ w3779 w3781 _ _ _ _ _ _ _ _ w3800 w3802 _]
          tunnel: w3373 -> [_ _ _ _ _ _ _ _ _ _ w3783 _ w3787 _ w3791 _ w3795 _ w3799 _ w3804]
          tunnel: w3372 -> [_ _ _ _ _ _ _ _ _ _ _ w3785 _ w3789 _ w3793 _ w3797 _ w3801 w3803]
          frame 0, Default {
          }
          frame 1 {
          }
          frame 2 {
          }
          frame 3 {
          }
          frame 4 {
          }
          frame 5 {
          }
          frame 6 {
          }
          frame 7 {
          }
          frame 8 {
          }
          frame 9 {
          }
          frame 10 {
          }
          frame 11 {
          }
          frame 12 {
          }
          frame 13 {
          }
          frame 14 {
          }
          frame 15 {
          }
          frame 16 {
          }
          frame 17 {
          }
          frame 18 {
          }
          frame 19 {
          }
          frame 20 {
          }
        }
        n1260 = case shown="19" "差分X2" {
          tunnel: w3377 -> [w3709 w3711 w3713 w3715 _ _ _ _ _ _ w3729 w3731 _ _ _ _ _ _ _ _ _]
          tunnel: w3376 -> [w3708 _ _ _ w3717 w3719 w3721 _ _ _ _ _ w3733 w3735 _ _ _ _ _ _ _]
          tunnel: w3368 -> [_ w3710 _ _ w3716 _ _ w3723 w3725 _ _ _ _ _ w3737 w3739 _ _ _ _ _]
          tunnel: w3375 -> [_ _ w3712 _ _ w3718 _ w3722 _ w3727 _ _ _ _ _ _ w3741 w3743 _ _ _]
          tunnel: [w3709 w3711 w3713 w3715 w3717 w3719 w3721 w3723 w3725 w3727 w3729 w3731 w3733 w3735 w3737 w3739 w3741 w3743 w3745 w3747 w3749] -> w3434
          tunnel: [w3708 w3710 w3712 w3714 w3716 w3718 w3720 w3722 w3724 w3726 w3728 w3730 w3732 w3734 w3736 w3738 w3740 w3742 w3744 w3746 w3748] -> w3438
          tunnel: w3374 -> [_ _ _ w3714 _ _ w3720 _ w3724 w3726 _ _ _ _ _ _ _ _ w3745 w3747 _]
          tunnel: w3373 -> [_ _ _ _ _ _ _ _ _ _ w3728 _ w3732 _ w3736 _ w3740 _ w3744 _ w3749]
          tunnel: w3372 -> [_ _ _ _ _ _ _ _ _ _ _ w3730 _ w3734 _ w3738 _ w3742 _ w3746 w3748]
          frame 0, Default {
          }
          frame 1 {
          }
          frame 2 {
          }
          frame 3 {
          }
          frame 4 {
          }
          frame 5 {
          }
          frame 6 {
          }
          frame 7 {
          }
          frame 8 {
          }
          frame 9 {
          }
          frame 10 {
          }
          frame 11 {
          }
          frame 12 {
          }
          frame 13 {
          }
          frame 14 {
          }
          frame 15 {
          }
          frame 16 {
          }
          frame 17 {
          }
          frame 18 {
          }
          frame 19 {
          }
          frame 20 {
          }
        }
        n1261 = case shown="19" "差分X3" {
          tunnel: w3377 -> [w3551 w3553 w3555 w3557 _ _ _ _ _ _ w3571 w3573 _ _ _ _ _ _ _ _ _]
          tunnel: w3376 -> [w3550 _ _ _ w3559 w3561 w3563 _ _ _ _ _ w3575 w3577 _ _ _ _ _ _ _]
          tunnel: w3368 -> [_ w3552 _ _ w3558 _ _ w3565 w3567 _ _ _ _ _ w3579 w3581 _ _ _ _ _]
          tunnel: w3375 -> [_ _ w3554 _ _ w3560 _ w3564 _ w3569 _ _ _ _ _ _ w3583 w3585 _ _ _]
          tunnel: [w3551 w3553 w3555 w3557 w3559 w3561 w3563 w3565 w3567 w3569 w3571 w3573 w3575 w3577 w3579 w3581 w3583 w3585 w3587 w3589 w3591] -> w3405
          tunnel: [w3550 w3552 w3554 w3556 w3558 w3560 w3562 w3564 w3566 w3568 w3570 w3572 w3574 w3576 w3578 w3580 w3582 w3584 w3586 w3588 w3590] -> w3401
          tunnel: w3374 -> [_ _ _ w3556 _ _ w3562 _ w3566 w3568 _ _ _ _ _ _ _ _ w3587 w3589 _]
          tunnel: w3373 -> [_ _ _ _ _ _ _ _ _ _ w3570 _ w3574 _ w3578 _ w3582 _ w3586 _ w3591]
          tunnel: w3372 -> [_ _ _ _ _ _ _ _ _ _ _ w3572 _ w3576 _ w3580 _ w3584 _ w3588 w3590]
          frame 0, Default {
          }
          frame 1 {
          }
          frame 2 {
          }
          frame 3 {
          }
          frame 4 {
          }
          frame 5 {
          }
          frame 6 {
          }
          frame 7 {
          }
          frame 8 {
          }
          frame 9 {
          }
          frame 10 {
          }
          frame 11 {
          }
          frame 12 {
          }
          frame 13 {
          }
          frame 14 {
          }
          frame 15 {
          }
          frame 16 {
          }
          frame 17 {
          }
          frame 18 {
          }
          frame 19 {
          }
          frame 20 {
          }
        }
        n1262 = case shown="19" "差分X" {
          tunnel: w3377 -> [w3819 w3821 w3823 w3825 _ _ _ _ _ _ w3839 w3841 _ _ _ _ _ _ _ _ _]
          tunnel: w3376 -> [w3818 _ _ _ w3827 w3829 w3831 _ _ _ _ _ w3843 w3845 _ _ _ _ _ _ _]
          tunnel: w3368 -> [_ w3820 _ _ w3826 _ _ w3833 w3835 _ _ _ _ _ w3847 w3849 _ _ _ _ _]
          tunnel: w3375 -> [_ _ w3822 _ _ w3828 _ w3832 _ w3837 _ _ _ _ _ _ w3851 w3853 _ _ _]
          tunnel: [w3819 w3821 w3823 w3825 w3827 w3829 w3831 w3833 w3835 w3837 w3839 w3841 w3843 w3845 w3847 w3849 w3851 w3853 w3855 w3857 w3859] -> w3455
          tunnel: [w3818 w3820 w3822 w3824 w3826 w3828 w3830 w3832 w3834 w3836 w3838 w3840 w3842 w3844 w3846 w3848 w3850 w3852 w3854 w3856 w3858] -> w3451
          tunnel: w3374 -> [_ _ _ w3824 _ _ w3830 _ w3834 w3836 _ _ _ _ _ _ _ _ w3855 w3857 _]
          tunnel: w3373 -> [_ _ _ _ _ _ _ _ _ _ w3838 _ w3842 _ w3846 _ w3850 _ w3854 _ w3859]
          tunnel: w3372 -> [_ _ _ _ _ _ _ _ _ _ _ w3840 _ w3844 _ w3848 _ w3852 _ w3856 w3858]
          frame 0, Default {
          }
          frame 1 {
          }
          frame 2 {
          }
          frame 3 {
          }
          frame 4 {
          }
          frame 5 {
          }
          frame 6 {
          }
          frame 7 {
          }
          frame 8 {
          }
          frame 9 {
          }
          frame 10 {
          }
          frame 11 {
          }
          frame 12 {
          }
          frame 13 {
          }
          frame 14 {
          }
          frame 15 {
          }
          frame 16 {
          }
          frame 17 {
          }
          frame 18 {
          }
          frame 19 {
          }
          frame 20 {
          }
        }
        n1263 = Index Array(array=w3443, index (row)="Y2") -> (element=w3444:dbl[])  [unwired: 1 in]
        n1264 = Index Array(array=w3396, index (row)="Y3") -> (element=w3395:dbl[])  [unwired: 1 in]
        n1265 = Index Array(array=w3446, index (row)="Y") -> (element=w3445:dbl[])  [unwired: 1 in]
        n1266 = Index Array(array=w3434, index (row)="X2") -> (element=w3433:dbl[])  [unwired: 1 in]
        n1267 = Index Array(array=w3405, index (row)="X3") -> (element=w3406:dbl[])  [unwired: 1 in]
        n1268 = Index Array(array=w3455, index (row)="X") -> (element=w3456:dbl[])  [unwired: 1 in]
        n1269 = Index Array(array=w3439, index (row)="Y2") -> (element=w3441:dbl[])  [unwired: 1 in]
        n1270 = Index Array(array=w3400, index (row)="Y3") -> (element=w3398:dbl[])  [unwired: 1 in]
        n1271 = Index Array(array=w3450, index (row)="Y") -> (element=w3448:dbl[])  [unwired: 1 in]
        n1272 = Index Array(array=w3438, index (row)="X2") -> (element=w3436:dbl[])  [unwired: 1 in]
        n1273 = Index Array(array=w3401, index (row)="X3") -> (element=w3403:dbl[])  [unwired: 1 in]
        n1274 = Index Array(array=w3451, index (row)="X") -> (element=w3453:dbl[])  [unwired: 1 in]
        n1275 = Delete From Array(array=w3444, length=w3382, index=w3371) -> (array with subset deleted=w3442:dbl[])  [unwired: 1 out]
        n1276 = Delete From Array(array=w3395, length=w3384, index=w3371) -> (array with subset deleted=w3397:dbl[])  [unwired: 1 out]
        n1277 = Delete From Array(array=w3445, length=w3380, index=w3371) -> (array with subset deleted=w3447:dbl[])  [unwired: 1 out]
        n1278 = Delete From Array(array=w3433, length=w3381, index=w3371) -> (array with subset deleted=w3435:dbl[])  [unwired: 1 out]
        n1279 = Delete From Array(array=w3406, length=w3383, index=w3371) -> (array with subset deleted=w3404:dbl[])  [unwired: 1 out]
        n1280 = Delete From Array(array=w3456, length=w3379, index=w3371) -> (array with subset deleted=w3454:dbl[])  [unwired: 1 out]
        n1281 = Delete From Array(array=w3441, length=w3382, index=w3371) -> (array with subset deleted=w3440:dbl[])  [unwired: 1 out]
        n1282 = Delete From Array(array=w3398, length=w3384, index=w3371) -> (array with subset deleted=w3399:dbl[])  [unwired: 1 out]
        n1283 = Delete From Array(array=w3448, length=w3380, index=w3371) -> (array with subset deleted=w3449:dbl[])  [unwired: 1 out]
        n1284 = Delete From Array(array=w3436, length=w3381, index=w3371) -> (array with subset deleted=w3437:dbl[])  [unwired: 1 out]
        n1285 = Delete From Array(array=w3403, length=w3383, index=w3371) -> (array with subset deleted=w3402:dbl[])  [unwired: 1 out]
        n1286 = Delete From Array(array=w3453, length=w3379, index=w3371) -> (array with subset deleted=w3452:dbl[])  [unwired: 1 out]
        n1287 = xnode "公式 Aa 4"("X1"=w3435, "X2"=w3437) -> ("结果"=w3413:dbl[])  [unwired: 1 in, 1 out]
        n1288 = xnode "公式 Aa 6"("X1"=w3404, "X2"=w3402) -> ("结果"=w3408:dbl[])  [unwired: 1 in, 1 out]
        n1289 = xnode "公式 Aa 5"("X1"=w3442, "X2"=w3440) -> ("结果"=w3411:dbl[])  [unwired: 1 in, 1 out]
        n1290 = xnode "公式 Aa 7"("X1"=w3397, "X2"=w3399) -> ("结果"=w3410:dbl[])  [unwired: 1 in, 1 out]
        n1291 = xnode "公式 Aa 3"("X1"=w3447, "X2"=w3449) -> ("结果"=w3416:dbl[])  [unwired: 1 in, 1 out]
        n1292 = xnode "公式 Aa 2"("X1"=w3454, "X2"=w3452) -> ("结果"=w3419:dbl[])  [unwired: 1 in, 1 out]
        n1293 = call "绘图-分段颜色-差分.vi"("分段颜色"=w3370, "基准索引"=w3369, "光谱值"=w3416, "清空"="波长差分B") -> ("数组"=w3415:dbl[][])  [unwired: 7 in]
        n1294 = call "绘图-分段颜色-差分.vi"("分段颜色"=w3370, "基准索引"=w3369, "光谱值"=w3413, "清空"="波长差分A2") -> ("数组"=w3414:dbl[][])  [unwired: 7 in]
        n1295 = call "绘图-分段颜色-差分.vi"("分段颜色"=w3370, "基准索引"=w3369, "光谱值"=w3408, "清空"="波长差分A3") -> ("数组"=w3407:dbl[][])  [unwired: 7 in]
        n1296 = call "绘图-分段颜色-差分.vi"("分段颜色"=w3370, "基准索引"=w3369, "光谱值"=w3411, "清空"="波长差分B2") -> ("数组"=w3412:dbl[][])  [unwired: 7 in]
        n1297 = call "绘图-分段颜色-差分.vi"("分段颜色"=w3370, "基准索引"=w3369, "光谱值"=w3410, "清空"="波长差分B3") -> ("数组"=w3409:dbl[][])  [unwired: 7 in]
        n1298 = call "绘图-分段颜色-差分.vi"("分段颜色"=w3370, "基准索引"=w3369, "光谱值"=w3419, "清空"="波长差分A") -> ("数组"=w3418:dbl[][])  [unwired: 7 in]
        n1299 = case shown="True" "波长差分B3" {
          selector: "波长差分B3" -> [_ w3459]
          frame False {
          }
          frame True {
            n1300 = Not(x=w3459) -> (.not. x?=w3458:bool)
            n1301 = local write "波长差分B3"(w3458) -> ()
          }
        }
        n1302 = case shown="True" "波长差分B" {
          selector: "波长差分B" -> [_ w3597]
          frame False {
          }
          frame True {
            n1303 = Not(x=w3597) -> (.not. x?=w3596:bool)
            n1304 = local write "波长差分B"(w3596) -> ()
          }
        }
        n1305 = case shown="True" "波长差分A" {
          selector: "波长差分A" -> [_ w3599]
          frame False {
          }
          frame True {
            n1306 = Not(x=w3599) -> (.not. x?=w3598:bool)
            n1307 = local write "波长差分A"(w3598) -> ()
          }
        }
        n1308 = case shown="True" "波长差分B2" {
          selector: "波长差分B2" -> [_ w3593]
          frame False {
          }
          frame True {
            n1309 = Not(x=w3593) -> (.not. x?=w3592:bool)
            n1310 = local write "波长差分B2"(w3592) -> ()
          }
        }
        n1311 = case shown="True" "波长差分A3" {
          selector: "波长差分A3" -> [_ w3461]
          frame False {
          }
          frame True {
            n1312 = Not(x=w3461) -> (.not. x?=w3460:bool)
            n1313 = local write "波长差分A3"(w3460) -> ()
          }
        }
        n1314 = case shown="True" "波长差分A2" {
          selector: "波长差分A2" -> [_ w3595]
          frame False {
          }
          frame True {
            n1315 = Not(x=w3595) -> (.not. x?=w3594:bool)
            n1316 = local write "波长差分A2"(w3594) -> ()
          }
        }
        n1317 = xnode "公式 2"("X1"=w3414, "X2"=w3412, "k"="k2") -> ("结果"=→"F_dAd_2":dbl[][])  [unwired: 1 in, 1 out]
        n1318 = xnode "公式 3"("X1"=w3407, "X2"=w3409, "k"="k3") -> ("结果"=→"F_dAd_3":dbl[][])  [unwired: 1 in, 1 out]
        n1319 = call <vilib>:"Add State(s) to Queue__jki_lib_state_machine.vi"("State(s) in (\"\")"=w3365) -> ("States Out"=w3366:string)  [unwired: 14 in]
        n1320 = xnode "公式"("X1"=w3418, "X2"=w3415, "k"="k") -> ("结果"=→"F_dAd_1":dbl[][])  [unwired: 1 in, 1 out]
      }
      frame "---------- Macro ----------" {
        # "#CSM \"Category Seperator\"\nDo not put any code in this frame."
        n1321 = call <vilib>:"Add State(s) to Queue__JKI_lib_State_Machine.vi"("State(s) in (\"\")"=w3862) -> ("States Out"=w3861:string)  [unwired: 14 in]
      }
      frame "Macro: Initialize" {
        w3865 = "Data: Initialize\nInitialize Core Data\nUI: Initialize\n\n//Permanent registrations\nAcquired Data@Acquisition - <1> >> Data: Update Indicators -><register>\nAcquired Data@Acquisition - <1> >> API: Log@Logging - <1> -><register>\nWait Count@Acquisition - <1> >> Time: Wait Count@<1>_Time -><register>\n\n//Error registrations\nError Occurred@Acquisition - <1> >> Error Handler -><register>\nError Occurred@Logging - <1> >> Error Handler -><register>\nError Occurred@<1>_Time >> Error Handler -><register>\n\n//Dynamic registrations\n// 订阅/取消订阅\n//Status@SourceModule >> API@TargetModule -><register as interrupt>\n//UrgentEvent @SourceModule >> API@TargetModule -><register as status>\n\n\n\n//Launch Acquisition Module\n"  # Data: Initialize Initialize Core Data UI: Initialize  //Permanent registrations Acquired Data@Acquisition - <1> >> Data: Update Indicators -><register> Acquired Data@Acquisition - <1> >> API: Log@Logging - <1> -><register> Wait Count@Acquisition - <1> >> Time: Wait Count@<1>_Time -><register>  //Error registrations Error Occurred@Acquisition - <1> >> Error Handler -><register> Error Occurred@Logging - <1> >> Error Handler -><register> Error Occurred@<1>_Time >> Error Handler -><register>  //Dynamic registrations // 订阅/取消订阅 //Status@SourceModule >> API@TargetModule -><register as interrupt> //UrgentEvent @SourceModule >> API@TargetModule -><register as status>    //Launch Acquisition Module
        # "#CSM \"Macro: Initialize\"\nInitialization Macro (This is called once, when the VI starts)"
        n1322 = call-poly <userlib>:"Build Message with Arguments++.vi"("States With Replace Token"=w3865, "<1>"=w3864) -> ("States"=w3863:string)  [unwired: 13 in]
        n1323 = call <vilib>:"Add State(s) to Queue__JKI_lib_State_Machine.vi"("State(s) in Front (\"\")"=w3863, "State(s) in (\"\")"=w3868) -> ("States Out"=w3867:string)  [unwired: 13 in]
      }
      frame "Macro: Start" {
        w3893 = "-" ("字符串")
        w3899 = 1  # 起始周期
        n1324 = Unbundle By Name(w3883) -> ("Time and Data.当前运行信息.当前周期"=w3900:i32, "Time and Data.当前运行信息.测量周期"=w3898:i32, "Sample Settings.CSM.CSM Name"=w3891:string)
        n1325 = call "Convert API String Arguments to Data.vim"("Reference Type"=FALSE, "API String"=w3897) -> ("Data"=w3895:bool)  [unwired: 6 in, 1 out]
        n1326 = Get Date/Time In Seconds() -> (seconds since 1Jan1904=w3878:timestamp)
        n1327 = Format Date/Time String(time format string (%c)="%Y%m%d-%H%M%S" ("时间格式字符串(%c)"), seconds (now)=w3878) -> (date/time string=w3890:string)  [unwired: 1 in]
        n1328 = case shown="\"5环-双测头\"" "测头类型" {
          tunnel: "信号采集设备和供电" -> [w3921 w3927 w3932 w3938 w3944]
          tunnel: [w3919 w3925 w3931 w3937 w3943] -> w3876
          tunnel: [w3918 TRUE w3930 w3936 TRUE] -> _
          tunnel: [w3918 FALSE w3930 w3936 FALSE] -> _
          tunnel: [u8 5 u8 5 u8 5 u8 7 u8 7] -> w3875
          frame "5环-单测头", Default {
            w3918 = FALSE
            n1329 = Concatenate Strings(w3921, "/ai1:5" ("字符串")) -> (w3919:string)
          }
          frame "5环-双测头" {
            n1330 = Concatenate Strings(w3927, "/ai1:7, " ("字符串"), w3927, "/ai16:18" ("字符串")) -> (w3925:string)
          }
          frame "5环-三测头" {
            w3930 = TRUE
            n1331 = Concatenate Strings(w3932, "/ai1:7, " ("字符串"), w3932, "/ai16:23" ("字符串")) -> (w3931:string)
          }
          frame "7环-单测头" {
            w3936 = FALSE
            n1332 = Concatenate Strings(w3938, "/ai1:7" ("字符串")) -> (w3937:string)
          }
          frame "7环-双测头" {
            n1333 = Concatenate Strings(w3944, "/ai1:7, " ("字符串"), w3944, "/ai16:20" ("字符串")) -> (w3943:string)
          }
        }
        n1334 = local read "校准模式"() -> (w3871:T5)
        n1335 = Not Equal?(x="数据文件前缀", y="") -> (x != y?=w3901:bool)
        n1336 = Concatenate Strings(w3890, w3893, w3891, w3893) -> (w3892:string)
        n1337 = To Byte Integer(number="测量波长") -> (8bit integer=w3869:i8[])
        n1338 = Compound Arithmetic op=AND ("复合运算")(w3901, w3895) -> (w3888:bool)
        n1339 = Select(t=w3900, s=w3888, f=w3899) -> (s? t:f=w3881:i32)
        n1340 = Select(t=w3898, s=w3888, f=w3899) -> (s? t:f=w3880:i32)
        n1341 = Select(t="数据文件前缀", s=w3888, f=w3892) -> (s? t:f=w3879:string)
        n1342 = local write "数据文件前缀"(w3879) -> ()
        n1343 = Build Array (concatenate)(i8 -1, w3869) -> (w3882:i8[])
        n1344 = in-place {
          in-place-border: "测量波长" -> [w3916]
          in-place-border: w3882 -> [w3915]
          in-place-border: w3871 -> [w3914]
          in-place-border: w3881 -> [w3913]
          in-place-border: w3880 -> [w3912]
          in-place-border: w3879 -> [w3911]
          in-place-border: w3878 -> [w3910]
          in-place-border: "信号采集设备和供电" -> [w3909]
          in-place-border: w3876 -> [w3908]
          in-place-border: w3875 -> [w3907]
          in-place-border: "测头类型" -> [w3906]
          n1345 = in-place-cluster #27(w3883) -> ()  [unwired: 11 out]
          n1346 = in-place-cluster #27("Indicators.控制.测量波长"=w3916, "Sample Settings.设备信息.初始索引子集"=w3915, "Sample Settings.校准.校准模式"=w3914, "Sample Settings.测量.起始周期"=w3913, "Sample Settings.测量.起始测量周期"=w3912, "Sample Settings.图表相关.文件-时间"=w3911, "Indicators.图表相关.程序开始时间"=w3910, "Indicators.控制.信号采集设备和供电"=w3909, "Sample Settings.设备信息.模拟信号采集通道"=w3908, "Sample Settings.设备信息.环数"=w3907, "Indicators.控制.测头类型"=w3906) -> (w3873:T20)
        }
        n1347 = Select(t="", s=w3888, f="Plot: Reset") -> (s? t:f=w3885:string)
        n1348 = call <vilib>:"Add State(s) to Queue__JKI_lib_State_Machine.vi"("State(s) in Front (\"\")"="UI Initialize Start" ("State(s) in Front (\"\")"), "State(s) in (\"\")"=w3885) -> ("States Out"=w3884:string)  [unwired: 13 in]
        n1349 = call <vilib>:"Add State(s) to Queue__JKI_lib_State_Machine.vi"("State(s) in Front (\"\")"=w3884, "State(s) in (\"\")"=w3905) -> ("States Out"=w3904:string)  [unwired: 13 in]
      }
      frame "Macro: Stop" {
        # "#CSM \"Macro: Exit\"\nExit Macro (This is called once, when the VI exits)"
        n1350 = property on="开始" class="Bool"("DisabledEnum"=T11."Enabled" ("禁用")) -> ()  [unwired: 2 in, 2 out]
        n1351 = call-poly <userlib>:"Build Message with Arguments++.vi"("States With Replace Token"="//Send Message to Other CSM Modules\nAPI: Stop -@ Acquisition - <1>\nAPI: Stop -@ Logging - <1>", "<1>"=w3949) -> ("States"=w3948:string)  [unwired: 13 in]
        n1352 = call <vilib>:"Add State(s) to Queue__JKI_lib_State_Machine.vi"("State(s) in Front (\"\")"=w3948, "State(s) in (\"\")"=w3953) -> ("States Out"=w3952:string)  [unwired: 13 in]
      }
      frame "Macro: Exit" {
        w3958 = "//Exit\nMacro: Exit-@Acquisition - <1>\nMacro: Exit-@Logging - <1>\nMacro: Exit-@<1>_Time\n\n//Permanent unregistrations\nAcquired Data@Acquisition - <1> >> Data: Update Indicators -><unregister>\nAcquired Data@Acquisition - <1> >> API: Log@Logging - <1> -><unregister>\nWait Count@Acquisition - <1> >> Time: Wait Count@<1>_Time -><unregister>\n\n//Permanent unregistrations\nError Occurred@Acquisition - <1> >> Error Handler -><unregister>\nError Occurred@Logging - <1> >> Error Handler -><unregister>\nError Occurred@<1>_Time >> Error Handler -><unregister>\n\nData: Cleanup\nExit"  # //Exit Macro: Exit-@Acquisition - <1> Macro: Exit-@Logging - <1> Macro: Exit-@<1>_Time  //Permanent unregistrations Acquired Data@Acquisition - <1> >> Data: Update Indicators -><unregister> Acquired Data@Acquisition - <1> >> API: Log@Logging - <1> -><unregister> Wait Count@Acquisition - <1> >> Time: Wait Count@<1>_Time -><unregister>  //Permanent unregistrations Error Occurred@Acquisition - <1> >> Error Handler -><unregister> Error Occurred@Logging - <1> >> Error Handler -><unregister> Error Occurred@<1>_Time >> Error Handler -><unregister>  Data: Cleanup Exit
        # "#CSM \"Macro: Exit\"\nExit Macro (This is called once, when the VI exits)"
        n1353 = disable-structure shown="禁用" {
          frame Disabled {
            # "#NOTE\nHelper VI is equivalent to other case"
            n1354 = call <userlib>:"CSM - Build Exit Messages of CSMs.vi"("State With Arguments (\"Macro: Exit“)"="Macro: Exit" ("State with Arguments(\"Macro: Exit“)"), "CSMs"=string[] ["AcquisitionTP1", "//LoggingTP1"]) -> ()  [unwired: 13 in, 1 out]
          }
          frame Enabled {
          }
        }
        n1355 = local write "程序状态"("已停止" ("程序状态")) -> ()
        n1356 = property on="开始" class="Bool"("DisabledEnum"=T11."Enabled" ("禁用")) -> ()  [unwired: 2 in, 2 out]
        n1357 = call-poly <userlib>:"Build Message with Arguments++.vi"("States With Replace Token"=w3958, "<1>"=w3957) -> ("States"=w3956:string)  [unwired: 13 in]
        n1358 = call <vilib>:"Add State(s) to Queue__JKI_lib_State_Machine.vi"("State(s) in Front (\"\")"=w3956, "State(s) in (\"\")"=w3961) -> ("States Out"=w3960:string)  [unwired: 13 in]
      }
      frame "Macro: Pause" {
      }
      frame "---------- Plot ----------" {
        # "#CSM \"Category Seperator\"\nDo not put any code in this frame."
        n1359 = call <vilib>:"Add State(s) to Queue__JKI_lib_State_Machine.vi"("State(s) in (\"\")"=w3967) -> ("States Out"=w3968:string)  [unwired: 14 in]
      }
      frame "Plot: Reset" {
        w3972 = TRUE
        # "#CSM \"Category Seperator\"\nDo not put any code in this frame."
        n1360 = local write "45AD"(dbl[][] []) -> ()
        n1361 = local write "时间-周期对照"(string[][] []) -> ()
        n1362 = property on="时间-周期" class="WFChart (严格)"("History Data"=waveform(i32)[] [] ("历史数据")) -> ()  [unwired: 2 in, 2 out]
        n1363 = local write "波长差分A"(w3972) -> ()
        n1364 = local write "波长差分B"(w3972) -> ()
        n1365 = local write "波长差分A2"(w3972) -> ()
        n1366 = local write "波长差分B2"(w3972) -> ()
        n1367 = local write "波长差分A3"(w3972) -> ()
        n1368 = local write "波长差分B3"(w3972) -> ()
        n1369 = local write "R单环Aa"(w3972) -> ()
        n1370 = local write "R单环Ab"(w3972) -> ()
        n1371 = local write "R单环Ac"(w3972) -> ()
        n1372 = local write "R单环Ba"(w3972) -> ()
        n1373 = local write "R单环Bb"(w3972) -> ()
        n1374 = local write "R单环Bc"(w3972) -> ()
        n1375 = local write "R单环Ca"(w3972) -> ()
        n1376 = local write "R单环Cb"(w3972) -> ()
        n1377 = local write "R单环Cc"(w3972) -> ()
        n1378 = local write "R差分Dc"(w3972) -> ()
        n1379 = local write "R差分Aa"(w3972) -> ()
        n1380 = local write "R差分Ab"(w3972) -> ()
        n1381 = local write "R差分Ac"(w3972) -> ()
        n1382 = local write "R差分Ba"(w3972) -> ()
        n1383 = local write "R差分Bb"(w3972) -> ()
        n1384 = local write "R差分Bc"(w3972) -> ()
        n1385 = local write "R差分Ca"(w3972) -> ()
        n1386 = local write "R差分Cb"(w3972) -> ()
        n1387 = local write "R差分Cc"(w3972) -> ()
        n1388 = local write "R差分Da"(w3972) -> ()
        n1389 = local write "R差分Db"(w3972) -> ()
        n1390 = call <vilib>:"Add State(s) to Queue__JKI_lib_State_Machine.vi"("State(s) in (\"\")"=w3974) -> ("States Out"=w3975:string)  [unwired: 14 in]
        n1391 = local write "R差分Ea"(w3972) -> ()
        n1392 = local write "R差分Ec"(w3972) -> ()
        n1393 = local write "R差分Fa"(w3972) -> ()
        n1394 = local write "R差分Fc"(w3972) -> ()
        n1395 = local write "R差分Gc"(w3972) -> ()
        n1396 = local write "R差分Hb"(w3972) -> ()
        n1397 = local write "R差分Hc"(w3972) -> ()
        n1398 = local write "R差分Eb"(w3972) -> ()
        n1399 = local write "R差分Fb"(w3972) -> ()
        n1400 = local write "R差分Ga"(w3972) -> ()
        n1401 = local write "R差分Gb"(w3972) -> ()
        n1402 = local write "R差分Ha"(w3972) -> ()
      }
      frame "Plot: sg_justify" {
        n1403 = control-ref of="F单环Aa"() -> (w3981:refnum<vi>)
        n1404 = control-ref of="F单环Ab"() -> (w3982:refnum<vi>)
        n1405 = control-ref of="F单环Ac"() -> (w3983:refnum<vi>)
        n1406 = control-ref of="F单环Ba"() -> (w3984:refnum<vi>)
        n1407 = control-ref of="F单环Bb"() -> (w3985:refnum<vi>)
        n1408 = control-ref of="F单环Bc"() -> (w3986:refnum<vi>)
        n1409 = control-ref of="F单环Ca"() -> (w3987:refnum<vi>)
        n1410 = control-ref of="F单环Cb"() -> (w3988:refnum<vi>)
        n1411 = control-ref of="F单环Cc"() -> (w3989:refnum<vi>)
        n1412 = call "Convert API String Arguments to Data.vim"("Reference Type"=T12 {"上限"=0.0, "下限"=0.0, "图范围"=enum."自动"} ("簇"), "API String"=w3979) -> ("Data"=w3991:T12)  [unwired: 6 in, 1 out]
        n1413 = Unbundle(w3991) -> ("上限"=w3993:dbl, "下限"=w3994:dbl, "图范围"=w3992:enum32{"自动", "固定", "自定义"})
        n1414 = Build Array(w3981, w3982, w3983, w3984, w3985, w3986, w3987, w3988, w3989) -> (w3990:refnum<vi>[])
        n1415 = case shown="\"固定\"" w3992 {
          tunnel: w3990 -> [w3997 w4000 w4005]
          tunnel: w3993 -> [_ _ w4004]
          tunnel: w3994 -> [_ _ w4003]
          frame "自动", Default {
            n1416 = for {
              tunnel: w3997 -> [w3998] mode=indexing
              n1417 = property class="WFGraph"(reference=w3998, "YScale.ScaleFit"=u8 2 ("Y标尺.标尺调节")) -> ()  [unwired: 1 in, 2 out]
            }
          }
          frame "固定" {
            n1418 = for {
              tunnel: w4000 -> [w4001] mode=indexing
              n1419 = property class="WFGraph"(reference=w4001, "YScale.ScaleFit"=u8 0 ("Y标尺.标尺调节")) -> ()  [unwired: 1 in, 2 out]
            }
          }
          frame "自定义" {
            n1420 = flat-sequence {
              tunnel: w4005 -> [w4006]
              tunnel: w4005 -> [w4012]
              tunnel: w4004 -> [w4011]
              tunnel: w4003 -> [w4010]
              frame #0 {
                n1421 = for {
                  tunnel: w4006 -> [w4007] mode=indexing
                  n1422 = property class="WFGraph"(reference=w4007, "YScale.ScaleFit"=u8 0 ("Y标尺.标尺调节")) -> ()  [unwired: 1 in, 2 out]
                }
              }
              frame #1 {
                n1423 = Wait (ms)(milliseconds to wait=u32 10 ("等待时间（毫秒）")) -> ()  [unwired: 1 out]
              }
              frame #2 {
                n1424 = for {
                  tunnel: w4011 -> [w4015]
                  tunnel: w4010 -> [w4014]
                  tunnel: w4012 -> [w4013] mode=indexing
                  n1425 = property class="WFGraph"(reference=w4013, "YScale.Maximum"=w4015, "YScale.Minimum"=w4014) -> ()  [unwired: 1 in, 2 out]
                }
              }
            }
          }
        }
        n1426 = call <vilib>:"Add State(s) to Queue__JKI_lib_State_Machine.vi"("State(s) in (\"\")"=w3977) -> ("States Out"=w3978:string)  [unwired: 14 in]
      }
      frame "Plot: diff_justify" {
        n1427 = control-ref of="F差分Aa"() -> (w4022:refnum<vi>)
        n1428 = control-ref of="F差分Ac"() -> (w4024:refnum<vi>)
        n1429 = control-ref of="F差分Bb"() -> (w4026:refnum<vi>)
        n1430 = control-ref of="F差分Ca"() -> (w4028:refnum<vi>)
        n1431 = control-ref of="F差分Cc"() -> (w4030:refnum<vi>)
        n1432 = control-ref of="F差分Db"() -> (w4032:refnum<vi>)
        n1433 = control-ref of="F差分Ea"() -> (w4034:refnum<vi>)
        n1434 = control-ref of="F差分Ec"() -> (w4036:refnum<vi>)
        n1435 = control-ref of="F差分Fb"() -> (w4038:refnum<vi>)
        n1436 = control-ref of="F差分Ga"() -> (w4040:refnum<vi>)
        n1437 = control-ref of="F差分Gc"() -> (w4042:refnum<vi>)
        n1438 = control-ref of="F差分Hb"() -> (w4044:refnum<vi>)
        n1439 = control-ref of="F_dAd_1"() -> (w4046:refnum<vi>)
        n1440 = control-ref of="F_dAd_3"() -> (w4048:refnum<vi>)
        n1441 = control-ref of="F差分Ab"() -> (w4023:refnum<vi>)
        n1442 = control-ref of="F差分Ba"() -> (w4025:refnum<vi>)
        n1443 = control-ref of="F差分Bc"() -> (w4027:refnum<vi>)
        n1444 = control-ref of="F差分Cb"() -> (w4029:refnum<vi>)
        n1445 = control-ref of="F差分Da"() -> (w4031:refnum<vi>)
        n1446 = control-ref of="F差分Dc"() -> (w4033:refnum<vi>)
        n1447 = control-ref of="F差分Eb"() -> (w4035:refnum<vi>)
        n1448 = control-ref of="F差分Fa"() -> (w4037:refnum<vi>)
        n1449 = control-ref of="F差分Fc"() -> (w4039:refnum<vi>)
        n1450 = control-ref of="F差分Gb"() -> (w4041:refnum<vi>)
        n1451 = control-ref of="F差分Ha"() -> (w4043:refnum<vi>)
        n1452 = control-ref of="F差分Hc"() -> (w4045:refnum<vi>)
        n1453 = control-ref of="F_dAd_2"() -> (w4047:refnum<vi>)
        n1454 = Build Array(w4022, w4023, w4024, w4025, w4026, w4027, w4028, w4029, w4030, w4031, w4032, w4033, w4034, w4035, w4036, w4037, w4038, w4039, w4040, w4041, w4042, w4043, w4044, w4045, w4046, w4047, w4048) -> (w4049:refnum<vi>[])
        n1455 = call "Convert API String Arguments to Data.vim"("Reference Type"=T12 {"上限"=0.0, "下限"=0.0, "图范围"=enum."自动"} ("簇"), "API String"=w4016) -> ("Data"=w4018:T12)  [unwired: 6 in, 1 out]
        n1456 = Unbundle(w4018) -> ("上限"=w4020:dbl, "下限"=w4021:dbl, "图范围"=w4019:enum32{"自动", "固定", "自定义"})
        n1457 = case shown="\"自定义\"" w4019 {
          tunnel: w4049 -> [w4054 w4057 w4062]
          tunnel: w4020 -> [_ _ w4061]
          tunnel: w4021 -> [_ _ w4060]
          frame "自动", Default {
            n1458 = for {
              tunnel: w4054 -> [w4055] mode=indexing
              n1459 = property class="WFGraph"(reference=w4055, "YScale.ScaleFit"=u8 2 ("Y标尺.标尺调节")) -> ()  [unwired: 1 in, 2 out]
            }
          }
          frame "固定" {
            n1460 = for {
              tunnel: w4057 -> [w4058] mode=indexing
              n1461 = property class="WFGraph"(reference=w4058, "YScale.ScaleFit"=u8 0 ("Y标尺.标尺调节")) -> ()  [unwired: 1 in, 2 out]
            }
          }
          frame "自定义" {
            n1462 = flat-sequence {
              tunnel: w4062 -> [w4063]
              tunnel: w4062 -> [w4069]
              tunnel: w4061 -> [w4068]
              tunnel: w4060 -> [w4067]
              frame #0 {
                n1463 = for {
                  tunnel: w4063 -> [w4064] mode=indexing
                  n1464 = property class="WFGraph"(reference=w4064, "YScale.ScaleFit"=u8 0 ("Y标尺.标尺调节")) -> ()  [unwired: 1 in, 2 out]
                }
              }
              frame #1 {
                n1465 = Wait (ms)(milliseconds to wait=u32 10 ("等待时间（毫秒）")) -> ()  [unwired: 1 out]
              }
              frame #2 {
                n1466 = for {
                  tunnel: w4068 -> [w4072]
                  tunnel: w4067 -> [w4071]
                  tunnel: w4069 -> [w4070] mode=indexing
                  n1467 = property class="WFGraph"(reference=w4070, "YScale.Maximum"=w4072, "YScale.Minimum"=w4071) -> ()  [unwired: 1 in, 2 out]
                }
              }
            }
          }
        }
        n1468 = call <vilib>:"Add State(s) to Queue__JKI_lib_State_Machine.vi"("State(s) in (\"\")"=w4050) -> ("States Out"=w4051:string)  [unwired: 14 in]
      }
      frame "Plot: Add Delta Curve" {
        n1469 = Unbundle By Name(w4074) -> ("Sample Settings.测量.每波长测量次数"=w4073:i32)
        n1470 = local read "F差分Aa"() -> (w4099:dbl[][])
        n1471 = local read "F差分Ba"() -> (w4098:dbl[][])
        n1472 = local read "F差分Ca"() -> (w4097:dbl[][])
        n1473 = local read "F差分Fa"() -> (w4094:dbl[][])
        n1474 = local read "F差分Da"() -> (w4096:dbl[][])
        n1475 = local read "F差分Ea"() -> (w4095:dbl[][])
        n1476 = Array Size(array=w4099) -> (size(s)=w4079:i32[])
        n1477 = Array Size(array=w4098) -> (size(s)=w4080:i32[])
        n1478 = Array Size(array=w4097) -> (size(s)=w4081:i32[])
        n1479 = Array Size(array=w4096) -> (size(s)=w4082:i32[])
        n1480 = Array Size(array=w4095) -> (size(s)=w4083:i32[])
        n1481 = Array Size(array=w4094) -> (size(s)=w4084:i32[])
        n1482 = Subtract(x=w4079, y=w4073) -> (x-y=w4078:i32[])
        n1483 = Subtract(x=w4080, y=w4073) -> ()  [unwired: 1 out]
        n1484 = local read "A | Ad\n基准周期"() -> (w4091:i32)
        n1485 = Subtract(x=w4081, y=w4073) -> ()  [unwired: 1 out]
        n1486 = Subtract(x=w4082, y=w4073) -> ()  [unwired: 1 out]
        n1487 = Subtract(x=w4083, y=w4073) -> ()  [unwired: 1 out]
        n1488 = Subtract(x=w4084, y=w4073) -> ()  [unwired: 1 out]
        n1489 = Index Array(array=w4099) -> (element=w4076:dbl[])  [unwired: 2 in]
        n1490 = Index Array(array=w4078) -> (element=w4077:i32)  [unwired: 1 in]
        n1491 = Greater Than 0?(x=w4091) -> (x > 0?=w4092:bool)
        n1492 = Array Subset(array=w4076, index=w4077, length=w4073) -> (w4075:dbl[])
        n1493 = Array Subset(array=w4098, length (row)=w4073) -> ()  [unwired: 3 in, 1 out]
        n1494 = Array Subset(array=w4097, length (row)=w4073) -> ()  [unwired: 3 in, 1 out]
        n1495 = Array Subset(array=w4096, length (row)=w4073) -> ()  [unwired: 3 in, 1 out]
        n1496 = Array Subset(array=w4095, length (row)=w4073) -> ()  [unwired: 3 in, 1 out]
        n1497 = Array Subset(array=w4094, length (row)=w4073) -> ()  [unwired: 3 in, 1 out]
        n1498 = call <vilib>:"Std Deviation and Variance.vi"("X"=w4075) -> ("mean"=w4090:dbl)  [unwired: 1 in, 2 out]
        n1499 = call <vilib>:"Std Deviation and Variance.vi"() -> ("mean"=w4089:dbl)  [unwired: 2 in, 2 out]
        n1500 = call <vilib>:"Std Deviation and Variance.vi"() -> ("mean"=w4088:dbl)  [unwired: 2 in, 2 out]
        n1501 = call <vilib>:"Std Deviation and Variance.vi"() -> ("mean"=w4087:dbl)  [unwired: 2 in, 2 out]
        n1502 = call <vilib>:"Std Deviation and Variance.vi"() -> ("mean"=w4086:dbl)  [unwired: 2 in, 2 out]
        n1503 = call <vilib>:"Std Deviation and Variance.vi"() -> ("mean"=w4085:dbl)  [unwired: 2 in, 2 out]
        n1504 = Build Array(w4090, w4089, w4088, w4087, w4086, w4085) -> (w4093:dbl[])
        n1505 = case shown="True" w4092 {
          tunnel: w4093 -> [_ w4114]
          frame False {
            "添加/删除状态" <- "未添加成功——\"A | Ad基准周期\"应大于0"
          }
          frame True {
            n1506 = feedback #28(dbl[][] []) -> (w4106:dbl[][])
            n1507 = for "For循环" {
              tunnel: w4106 -> [w4124] mode=indexing
              tunnel: w4114 -> [w4123]
              tunnel: [w4121] -> w4105 mode=indexing
              n1508 = Equal?(x=w4124, y=w4123) -> (x = y?=w4122:bool[])
              n1509 = And Array Elements(Boolean array=w4122) -> (logical AND=w4121:bool)
            }
            n1510 = Or Array Elements(Boolean array=w4105) -> (logical OR=w4104:bool)
            n1511 = case shown="False" w4104 {
              tunnel: [w4118 w4120] -> w4108
              tunnel: w4106 -> [w4117 w4120]
              tunnel: w4114 -> [w4116 _]
              frame False {
                n1512 = Build Array (concatenate)(w4117, w4116) -> (w4118:dbl[][])
                n1513 = local write "添加/删除状态"("添加成功" ("添加状态")) -> ()
              }
              frame True {
                n1514 = local write "添加/删除状态"("请勿添加重复数据" ("添加状态")) -> ()
              }
            }
            n1515 = feedback-in #28(w4108) -> ()
            n1516 = Array Size(array=w4108) -> (size(s)=w4109:i32[])
            n1517 = Index Array(array=w4109) -> (element=w4110:i32)  [unwired: 1 in]
            n1518 = Subtract(x=w4110, y="显示数目") -> (x-y=w4111:i32)
            n1519 = Array Subset(array=w4108, index (row)=w4111, length (row)="显示数目") -> (→"45AD":dbl[][])  [unwired: 2 in]
          }
        }
        n1520 = call <vilib>:"Add State(s) to Queue__JKI_lib_State_Machine.vi"("State(s) in (\"\")"=w4100) -> ("States Out"=w4101:string)  [unwired: 14 in]
      }
      frame "Plot: Delete Delta Curve" {
        n1521 = local read "45AD"() -> (w4126:dbl[][])
        n1522 = Array Size(array=w4126) -> (size(s)=w4125:i32[])
        n1523 = Index Array(array=w4125) -> (element=w4127:i32)  [unwired: 1 in]
        n1524 = Greater?(x=w4127, y="删除项(按曲线编号)") -> (0:w4129:bool)
        n1525 = case shown="True" w4129 {
          tunnel: w4126 -> [_ w4137]
          tunnel: "删除项(按曲线编号)" -> [_ w4136]
          frame False {
            n1526 = local write "添加/删除状态"("删除失败，删除项过大。" ("添加状态")) -> ()
          }
          frame True {
            n1527 = Delete From Array(array=w4137, index (row)=w4136) -> (array with subset deleted=w4138:dbl[][])  [unwired: 2 in, 1 out]
            n1528 = local write "45AD"(w4138) -> ()
            n1529 = local write "添加/删除状态"("删除成功" ("添加状态")) -> ()
          }
        }
        n1530 = call <vilib>:"Add State(s) to Queue__JKI_lib_State_Machine.vi"("State(s) in (\"\")"=w4130) -> ("States Out"=w4131:string)  [unwired: 14 in]
      }
      frame "Plot: Set Base Cycle to Current" {
        # "以所设基准周期的最后一个点为基准\n\n0意为不设置基准周期，无论每波长测量几个点\n小于0意为不设置基准周期，无论每波长测量几个点\n大于0意为设置基准周期，无论每波长测量几个点"
        n1531 = Unbundle By Name(w4140) -> ("Sample Settings.测量.每波长测量次数"=w4144:i32, "Time and Data.当前运行信息.测量周期"=w4143:i32)
        n1532 = Decrement(x=w4143) -> (x-1=w4141:i32)
        n1533 = Multiply(x=w4144, y=w4141) -> (x*y=w4145:i32)
        n1534 = local write "A | Ad\n基准周期"(w4141) -> ()
        n1535 = Decrement(x=w4145) -> (x-1=w4142:i32)
        n1536 = in-place {
          in-place-border: w4142 -> [w4149]
          n1537 = in-place-cluster #29(w4140) -> ()  [unwired: 1 out]
          n1538 = in-place-cluster #29("Indicators.图表相关.基准索引"=w4149) -> (w4139:T20)
        }
        n1539 = call <vilib>:"Add State(s) to Queue__JKI_lib_State_Machine.vi"("State(s) in (\"\")"=w4146) -> ("States Out"=w4147:string)  [unwired: 14 in]
      }
      frame "Plot: Base Cycle Change" {
        # "以所设基准周期的最后一个点为基准\n\n0意为不设置基准周期，无论每波长测量几个点\n小于0意为不设置基准周期，无论每波长测量几个点\n大于0意为设置基准周期，无论每波长测量几个点"
        n1540 = call "Convert API String Arguments to Data.vim"("Reference Type"=1 ("A | Ad\n基准周期"), "API String"=w4155) -> ("Data"=w4150:i32)  [unwired: 6 in, 1 out]
        n1541 = Unbundle By Name(w4152) -> ("Sample Settings.测量.每波长测量次数"=w4157:i32, "Time and Data.当前运行信息.测量周期"=w4156:i32)
        n1542 = local write "A | Ad\n基准周期"(w4150) -> ()
        n1543 = Decrement(x=w4156) -> (x-1=w4159:i32)
        n1544 = Max & Min(x=w4150, y=w4159) -> (min(x,y)=w4160:i32)  [unwired: 1 out]
        n1545 = Multiply(x=w4157, y=w4160) -> (x*y=w4158:i32)
        n1546 = Decrement(x=w4158) -> (x-1=w4153:i32)
        n1547 = in-place {
          in-place-border: w4153 -> [w4164]
          n1548 = in-place-cluster #30(w4152) -> ()  [unwired: 1 out]
          n1549 = in-place-cluster #30("Indicators.图表相关.基准索引"=w4164) -> (w4151:T20)
        }
        n1550 = call <vilib>:"Add State(s) to Queue__JKI_lib_State_Machine.vi"("State(s) in (\"\")"=w4161) -> ("States Out"=w4162:string)  [unwired: 14 in]
      }
      frame "Plot: Temp Calib Set to 0" {
        n1551 = Unbundle By Name(w4166) -> ("Sample Settings.设备信息.环数"=w4169:u8)
        n1552 = call <vilib>:"Permute.vi"("k"=u32 2, "n"=w4169) -> ("nPk"=w4171:dbl)
        n1553 = Divide(x=w4171, y=2.0) -> (x/y=w4168:dbl)
        n1554 = Initialize Array(0.0 ("元素"), w4168, 6 ("维数大小")) -> (w4167:dbl[][])
        n1555 = local write "温度校准值（每度）"(w4167) -> ()
        n1556 = in-place {
          in-place-border: w4167 -> [w4178]
          n1557 = in-place-cluster #31(w4166) -> ()  [unwired: 1 out]
          n1558 = in-place-cluster #31("Indicators.校准.温度校准值（每度）"=w4178) -> (w4165:T20)
        }
        n1559 = call <vilib>:"Add State(s) to Queue__JKI_lib_State_Machine.vi"("State(s) in (\"\")"=w4175) -> ("States Out"=w4176:string)  [unwired: 14 in]
      }
      frame "Plot: Temp Calib Change" {
        n1560 = call "Convert API String Arguments to Data.vim"("Reference Type"=dbl[][] [[0.0, 0.0, 0.0, 0.0, 0.0, 0.0, 0.00013, 0.00013, 0.00013, 0.00013, 0.00013, 0.00013], [0.0, 0.0, 0.0, 0.0, 0.0, 0.0, 0.00013, 0.00013, 0.00013, 0.00013, 0.00013, 0.00013], [0.0, 0.0, 0.0, 0.0, 0.0, 0.0, 0.00013, 0.00013, 0.00013, 0.00013, 0.00013, 0.00013], [0.0, 0.0, 0.0, 0.0, 0.0, 0.0, 0.00013, 0.00013, 0.00013, 0.00013, 0.00013, 0.00013], [0.0, 0.0, 0.0, 0.0, 0.0, 0.0, 0.00013, 0.00013, 0.00013, 0.00013, 0.00013, 0.00013], [0.0, 0.0, 0.0, 0.0, 0.0, 0.0, 0.00013, 0.00013, 0.00013, 0.00013, 0.00013, 0.00013], [0.0, 0.0, 0.0, 0.0, 0.0, 0.0, 0.00013, 0.00013, 0.00013, 0.00013, 0.00013, 0.00013], [0.0, 0.0, 0.0, 0.0, 0.0, 0.0, 0.00013, 0.00013, 0.00013, 0.00013, 0.00013, 0.00013], [0.0, 0.0, 0.0, 0.0, 0.0, 0.0, 0.00013, 0.00013, 0.00013, 0.00013, 0.00013, 0.00013], [0.0, 0.0, 0.0, 0.0, 0.0, 0.0, 0.00013, 0.00013, 0.00013, 0.00013, 0.00013, 0.00013], [0.00013, 0.00013, 0.00013, 0.00013, 0.00013, 0.00013, 0.00013, 0.00013, 0.00013, 0.00013, 0.00013, 0.00013], [0.00013, 0.00013, 0.00013, 0.00013, 0.00013, 0.00013, 0.00013, 0.00013, 0.00013, 0.00013, 0.00013, 0.00013], [0.00013, 0.00013, 0.00013, 0.00013, 0.00013, 0.00013, 0.00013, 0.00013, 0.00013, 0.00013, 0.00013, 0.00013], [0.00013, 0.00013, 0.00013, 0.00013, 0.00013, 0.00013, 0.00013, 0.00013, 0.00013, 0.00013, 0.00013, 0.00013], [0.00013, 0.00013, 0.00013, 0.00013, 0.00013, 0.00013, 0.00013, 0.00013, 0.00013, 0.00013, 0.00013, 0.00013], [0.00013, 0.00013, 0.00013, 0.00013, 0.00013, 0.00013, 0.00013, 0.00013, 0.00013, 0.00013, 0.00013, 0.00013], [0.00013, 0.00013, 0.00013, 0.00013, 0.00013, 0.00013, 0.00013, 0.00013, 0.00013, 0.00013, 0.00013, 0.00013], [0.00013, 0.00013, 0.00013, 0.00013, 0.00013, 0.00013, 0.00013, 0.00013, 0.00013, 0.00013, 0.00013, 0.00013], [0.00013, 0.00013, 0.00013, 0.00013, 0.00013, 0.00013, 0.00013, 0.00013, 0.00013, 0.00013, 0.00013, 0.00013], [0.00013, 0.00013, 0.00013, 0.00013, 0.00013, 0.00013, 0.00013, 0.00013, 0.00013, 0.00013, 0.00013, 0.00013]] ("温度校准值（每度）"), "API String"=w4183) -> ("Data"=w4180:dbl[][])  [unwired: 6 in, 1 out]
        n1561 = in-place {
          in-place-border: w4180 -> [w4187]
          n1562 = in-place-cluster #32(w4181) -> ()  [unwired: 1 out]
          n1563 = in-place-cluster #32("Indicators.校准.温度校准值（每度）"=w4187) -> (w4179:T20)
        }
        n1564 = call <vilib>:"Add State(s) to Queue__JKI_lib_State_Machine.vi"("State(s) in (\"\")"=w4184) -> ("States Out"=w4185:string)  [unwired: 14 in]
      }
      frame "---------- API ----------" {
        # "#CSM \"Category Seperator\"\nDo not put any code in this frame."
        n1565 = call <vilib>:"Add State(s) to Queue__JKI_lib_State_Machine.vi"("State(s) in (\"\")"=w4188) -> ("States Out"=w4189:string)  [unwired: 14 in]
      }
      frame "API: Probe Up True" {
        n1566 = Unbundle By Name(w4192) -> ("Sample Settings.测量控制.测头拿起"=w4193:bool)
        n1567 = Wait (ms)(milliseconds to wait=u32 20 ("等待时间（毫秒）")) -> ()  [unwired: 1 out]
        n1568 = case shown="False" w4193 {
          tunnel: w4197 -> [w4217 _]
          tunnel: w4192 -> [w4200 w4221]
          tunnel: [w4201 w4221] -> w4196
          tunnel: w4195 -> [w4215 _]
          tunnel: [w4213 "" ("States Out")] -> w4194
          frame False {
            w4203 = TRUE ("测头供电")
            n1569 = call "Convert Data To API String Arguments.vim"("Data"=w4203) -> ("API String"=w4206:string)  [unwired: 7 in, 1 out]
            n1570 = local write "测头拿取"(w4203) -> ()
            n1571 = Not(x=w4203) -> (.not. x?=w4211:bool)
            n1572 = local read "计时方式"() -> (w4204:bool)
            n1573 = call "Convert Data To API String Arguments.vim"("Data"=w4211) -> ("API String"=w4205:string)  [unwired: 7 in, 1 out]
            n1574 = Concatenate Strings(w4215, " >> <param> -@ Acquisition - <1>" ("State")) -> (w4216:string)
            n1575 = case shown="True" w4204 {
              frame False {
              }
              frame True {
                n1576 = local write "开始/清零"(TRUE ("暂停/继续")) -> ()
              }
            }
            n1577 = call-poly <userlib>:"Build Message with Arguments++.vi"("States With Replace Token"=w4216, "<param>"=w4206, "<1>"=w4217) -> ("States"=w4210:string)  [unwired: 12 in]
            n1578 = call <vilib>:"Build State String with Arguments__JKI_lib_State_Machine.vi"("Arguments (\"\")"=w4205, "State"="API: Data Save") -> ("State with Arguments"=w4207:string)  [unwired: 4 in]
            n1579 = call <vilib>:"Build State String with Arguments__JKI_lib_State_Machine.vi"("Arguments (\"\")"=w4205, "State"="API: Probe Light") -> ("State with Arguments"=w4209:string)  [unwired: 4 in]
            n1580 = call <vilib>:"Add State(s) to Queue__jki_lib_state_machine.vi"("State(s) in Front (\"\")"=w4210, "State(s) in (\"\")"=w4207, "State(s) at Back (\"\")"=w4209) -> ("States Out"=w4213:string)  [unwired: 12 in]
            n1581 = in-place {
              in-place-border: Save_Delay."拿起" ("Indicators.Save Delay.进度") -> [w4219]
              in-place-border: w4203 -> [w4218]
              n1582 = in-place-cluster #33(w4200) -> ()  [unwired: 2 out]
              n1583 = in-place-cluster #33("Sample Settings.测量控制.测头拿起"=w4218, "Indicators.Save Delay.进度"=w4219) -> (w4201:T20)
            }
          }
          frame True {
          }
        }
        n1584 = call <vilib>:"Add State(s) to Queue__JKI_lib_State_Machine.vi"("State(s) in Front (\"\")"=w4194, "State(s) in (\"\")"=w4198) -> ("States Out"=w4199:string)  [unwired: 13 in]
      }
      frame "API: Probe Up False_Fast" {
        n1585 = Unbundle By Name(w4224) -> ("Sample Settings.测量控制.测头拿起"=w4223:bool)
        n1586 = case shown="True" w4223 {
          tunnel: w4228 -> [_ w4248]
          tunnel: w4224 -> [w4231 w4233]
          tunnel: [w4231 w4234] -> w4227
          tunnel: w4226 -> [_ w4247]
          tunnel: ["" ("States Out") w4238] -> w4225
          frame False {
          }
          frame True {
            w4236 = FALSE ("测头供电")
            n1587 = call "Convert Data To API String Arguments.vim"("Data"=w4236) -> ("API String"=w4242:string)  [unwired: 7 in, 1 out]
            n1588 = local write "测头拿取"(w4236) -> ()
            n1589 = Not(x=w4236) -> (.not. x?=w4243:bool)
            n1590 = call "Convert Data To API String Arguments.vim"("Data"=w4243) -> ("API String"=w4241:string)  [unwired: 7 in, 1 out]
            n1591 = Concatenate Strings(w4247, " >> <param> -@ Acquisition - <1>" ("State")) -> (w4246:string)
            n1592 = local read "计时方式"() -> (w4237:bool)
            n1593 = call-poly <userlib>:"Build Message with Arguments++.vi"("States With Replace Token"=w4246, "<param>"=w4242, "<1>"=w4248) -> ("States"=w4239:string)  [unwired: 12 in]
            n1594 = case shown="True" w4237 {
              frame False {
              }
              frame True {
                n1595 = local write "开始/清零"(TRUE ("暂停/继续")) -> ()
              }
            }
            n1596 = call <vilib>:"Build State String with Arguments__JKI_lib_State_Machine.vi"("Arguments (\"\")"=w4241, "State"="API: Probe Light") -> ("State with Arguments"=w4240:string)  [unwired: 4 in]
            n1597 = call <vilib>:"Add State(s) to Queue__jki_lib_state_machine.vi"("State(s) in Front (\"\")"=w4240, "State(s) in (\"\")"=w4239) -> ("States Out"=w4238:string)  [unwired: 13 in]
            n1598 = in-place {
              in-place-border: Save_Delay."Idle" ("Indicators.Save Delay.进度") -> [w4250]
              in-place-border: w4236 -> [w4249]
              n1599 = in-place-cluster #34(w4233) -> ()  [unwired: 2 out]
              n1600 = in-place-cluster #34("Sample Settings.测量控制.测头拿起"=w4249, "Indicators.Save Delay.进度"=w4250) -> (w4234:T20)
            }
          }
        }
        n1601 = call <vilib>:"Add State(s) to Queue__JKI_lib_State_Machine.vi"("State(s) in Front (\"\")"=w4225, "State(s) in (\"\")"=w4229) -> ("States Out"=w4230:string)  [unwired: 13 in]
      }
      frame "API: Probe Up False" {
        n1602 = Unbundle By Name(w4254) -> ("Sample Settings.测量控制.测头拿起"=w4252:bool, "Time and Data.当前运行信息.当前周期"=w4253:i32)
        n1603 = case shown="True" w4252 {
          tunnel: w4258 -> [_ w4280]
          tunnel: w4257 -> [_ w4267]
          tunnel: ["" ("States Out") w4279] -> w4256
          tunnel: [w4262 w4265] -> w4255
          tunnel: w4254 -> [w4262 w4266]
          tunnel: w4253 -> [_ w4263]
          frame False {
          }
          frame True {
            w4274 = FALSE ("测头供电")
            n1604 = Not(x=w4274) -> (.not. x?=w4277:bool)
            n1605 = call "Convert Data To API String Arguments.vim"("Data"=w4274) -> ("API String"=w4273:string)  [unwired: 7 in, 1 out]
            n1606 = call "Convert Data To API String Arguments.vim"("Data"=w4277) -> ("API String"=w4275:string)  [unwired: 7 in, 1 out]
            n1607 = local write "测头拿取"(w4274) -> ()
            n1608 = Concatenate Strings(w4267, " >> <param> -@ Acquisition - <1>" ("State")) -> (w4268:string)
            n1609 = Wait (ms)(milliseconds to wait=u32 20 ("等待时间（毫秒）")) -> ()  [unwired: 1 out]
            n1610 = call-poly <userlib>:"Build Message with Arguments++.vi"("States With Replace Token"=w4268, "<param>"=w4273, "<1>"=w4280) -> ("States"=w4276:string)  [unwired: 12 in]
            n1611 = call <vilib>:"Build State String with Arguments__JKI_lib_State_Machine.vi"("Arguments (\"\")"=w4275, "State"="API: Probe Light") -> ("State with Arguments"=w4272:string)  [unwired: 4 in]
            n1612 = call <vilib>:"Add State(s) to Queue__jki_lib_state_machine.vi"("State(s) in Front (\"\")"=w4276, "State(s) in (\"\")"=w4272, "State(s) at Back (\"\")"="API: Probe Up False_Disp") -> ("States Out"=w4279:string)  [unwired: 12 in]
            n1613 = in-place {
              in-place-border: w4263 -> [w4282]
              in-place-border: Save_Delay."放下-出光" ("Indicators.Save Delay.进度") -> [w4281]
              n1614 = in-place-cluster #35(w4266) -> ()  [unwired: 2 out]
              n1615 = in-place-cluster #35("Indicators.Save Delay.进度"=w4281, "Indicators.Save Delay.放下周期"=w4282) -> (w4265:T20)
            }
          }
        }
        n1616 = call <vilib>:"Add State(s) to Queue__JKI_lib_State_Machine.vi"("State(s) in Front (\"\")"=w4256, "State(s) in (\"\")"=w4259) -> ("States Out"=w4260:string)  [unwired: 13 in]
      }
      frame "API: Probe Up False_Disp" {
        n1617 = Unbundle By Name(w4287) -> ("Time and Data.Logging Settings.波长结束？"=w4283:bool, "Indicators.Save Delay.进度"=w4286:T13)
        n1618 = Wait (ms)(milliseconds to wait=u32 20 ("等待时间（毫秒）")) -> ()  [unwired: 1 out]
        n1619 = Equal?(x=Save_Delay."放下-出光", y=w4286) -> (x = y?=w4284:bool)
        n1620 = case shown="True" w4284 {
          tunnel: [w4293 w4295] -> w4290
          tunnel: w4287 -> [w4293 w4296]
          tunnel: ["" ("States Out") w4299] -> w4285
          tunnel: w4283 -> [_ _]
          frame False {
          }
          frame True {
            n1621 = in-place {
              in-place-border: Save_Delay."放下-显示" ("Indicators.Save Delay.进度") -> [w4300]
              n1622 = in-place-cluster #36(w4296) -> ()  [unwired: 1 out]
              n1623 = in-place-cluster #36("Indicators.Save Delay.进度"=w4300) -> (w4295:T20)
            }
            n1624 = call <vilib>:"Add State(s) to Queue__jki_lib_state_machine.vi"("State(s) in (\"\")"="API: Probe Up False_Save") -> ("States Out"=w4299:string)  [unwired: 14 in]
          }
        }
        n1625 = call <vilib>:"Add State(s) to Queue__JKI_lib_State_Machine.vi"("State(s) in (\"\")"=w4291, "State(s) at Back (\"\")"=w4285) -> ("States Out"=w4292:string)  [unwired: 13 in]
      }
      frame "API: Probe Up False_Save" {
        w4307 = Save_Delay."放下-显示" ("x")
        n1626 = Unbundle By Name(w4304) -> ("Sample Settings.测量控制.测头拿起"=w4305:bool, "Indicators.Save Delay.放下周期"=w4312:i32, "Time and Data.当前运行信息.当前周期"=w4311:i32, "Indicators.Save Delay.进度"=w4310:T13)
        n1627 = Less?(x=w4312, y=w4311) -> (x < y?=w4308:bool)
        n1628 = Equal?(x=w4310, y=w4307) -> (x = y?=w4306:bool)
        n1629 = case shown="True" w4306 {
          tunnel: ["" ("f") w4326] -> w4309
          tunnel: w4308 -> [_ w4322]
          tunnel: w4307 -> [w4320 w4325]
          tunnel: [w4320 w4324] -> w4303
          tunnel: [w4318 w4323] -> w4301
          tunnel: w4305 -> [w4318 w4321]
          frame False {
          }
          frame True {
            n1630 = case shown="True" w4322 {
              tunnel: ["API: Probe Up False_Save" w4336] -> w4326
              tunnel: w4325 -> [w4328 _]
              tunnel: [w4328 Save_Delay."Idle" ("Indicators.Save Delay.进度")] -> w4324
              tunnel: [w4327 FALSE ("Sample Settings.测量控制.测头拿起")] -> w4323
              tunnel: w4321 -> [w4327 _]
              frame False {
              }
              frame True {
                n1631 = local read "计时方式"() -> (w4331:bool)
                n1632 = call "Convert Data To API String Arguments.vim"("Data"=TRUE ("Sample Settings.测量控制.测头拿起")) -> ("API String"=w4334:string)  [unwired: 7 in, 1 out]
                n1633 = case shown="True" w4331 {
                  frame False {
                  }
                  frame True {
                    n1634 = local write "开始/清零"(TRUE ("暂停/继续")) -> ()
                  }
                }
                n1635 = call <vilib>:"Build State String with Arguments__JKI_lib_State_Machine.vi"("Arguments (\"\")"=w4334, "State"="API: Data Save") -> ("State with Arguments"=w4336:string)  [unwired: 4 in]
              }
            }
          }
        }
        n1636 = Wait (ms)(milliseconds to wait=u32 50 ("等待时间（毫秒）")) -> ()  [unwired: 1 out]
        n1637 = call <vilib>:"Add State(s) to Queue__JKI_lib_State_Machine.vi"("State(s) in (\"\")"=w4314, "State(s) at Back (\"\")"=w4309) -> ("States Out"=w4315:string)  [unwired: 13 in]
        n1638 = in-place {
          in-place-border: w4303 -> [w4317]
          in-place-border: w4301 -> [w4316]
          n1639 = in-place-cluster #37(w4304) -> ()  [unwired: 2 out]
          n1640 = in-place-cluster #37("Sample Settings.测量控制.测头拿起"=w4316, "Indicators.Save Delay.进度"=w4317) -> (w4302:T20)
        }
      }
      frame "API: Probe Power" {
        n1641 = call "Convert API String Arguments to Data.vim"("Reference Type"=TRUE ("测头供电"), "API String"=w4344) -> ("Data"=w4340:bool)  [unwired: 6 in, 1 out]
        n1642 = local write "测头供电"(w4340) -> ()
        n1643 = Concatenate Strings(w4342, " >> <param> -@ Acquisition - <1>" ("State")) -> (w4343:string)
        n1644 = call-poly <userlib>:"Build Message with Arguments++.vi"("States With Replace Token"=w4343, "<param>"=w4344, "<1>"=w4346) -> ("States"=w4345:string)  [unwired: 12 in]
        n1645 = in-place {
          in-place-border: w4340 -> [w4350]
          n1646 = in-place-cluster #38(w4339) -> ()  [unwired: 1 out]
          n1647 = in-place-cluster #38("Sample Settings.测量控制.测头供电"=w4350) -> (w4338:T20)
        }
        n1648 = call <vilib>:"Add State(s) to Queue__JKI_lib_State_Machine.vi"("State(s) in Front (\"\")"=w4345, "State(s) in (\"\")"=w4348) -> ("States Out"=w4349:string)  [unwired: 13 in]
      }
      frame "API: Probe Light" {
        n1649 = call "Convert API String Arguments to Data.vim"("Reference Type"=TRUE ("测头供电"), "API String"=w4357) -> ("Data"=w4352:bool)  [unwired: 6 in, 1 out]
        n1650 = local write "测头出光"(w4352) -> ()
        n1651 = Concatenate Strings(w4355, " >> <param> -@ Acquisition - <1>" ("State")) -> (w4354:string)
        n1652 = call-poly <userlib>:"Build Message with Arguments++.vi"("States With Replace Token"=w4354, "<param>"=w4357, "<1>"=w4359) -> ("States"=w4358:string)  [unwired: 12 in]
        n1653 = in-place {
          in-place-border: w4352 -> [w4363]
          n1654 = in-place-cluster #39(w4353) -> ()  [unwired: 1 out]
          n1655 = in-place-cluster #39("Sample Settings.测量控制.测头出光"=w4363) -> (w4351:T20)
        }
        n1656 = call <vilib>:"Add State(s) to Queue__JKI_lib_State_Machine.vi"("State(s) in Front (\"\")"=w4358, "State(s) in (\"\")"=w4361) -> ("States Out"=w4362:string)  [unwired: 13 in]
      }
      frame "API: Data Save" {
        n1657 = call "Convert API String Arguments to Data.vim"("Reference Type"=TRUE ("测头供电"), "API String"=w4370) -> ("Data"=w4365:bool)  [unwired: 6 in, 1 out]
        n1658 = local write "是否保存"(w4365) -> ()
        n1659 = Concatenate Strings(w4368, " >> <param> -@ Acquisition - <1>" ("State")) -> (w4367:string)
        n1660 = call-poly <userlib>:"Build Message with Arguments++.vi"("States With Replace Token"=w4367, "<param>"=w4370, "<1>"=w4372) -> ("States"=w4371:string)  [unwired: 12 in]
        n1661 = in-place {
          in-place-border: w4365 -> [w4376]
          n1662 = in-place-cluster #40(w4366) -> ()  [unwired: 1 out]
          n1663 = in-place-cluster #40("Sample Settings.测量控制.起始保存"=w4376) -> (w4364:T20)
        }
        n1664 = call <vilib>:"Add State(s) to Queue__JKI_lib_State_Machine.vi"("State(s) in Front (\"\")"=w4371, "State(s) in (\"\")"=w4374) -> ("States Out"=w4375:string)  [unwired: 13 in]
      }
      frame "API: Dark Curnt Mode" {
        n1665 = call "Convert API String Arguments to Data.vim"("Reference Type"=暗电流校准模式."逐周期" ("Sample Settings.校准.校准模式"), "API String"=w4384) -> ("Data"=w4379:T5)  [unwired: 6 in, 1 out]
        n1666 = Concatenate Strings(w4382, " >> <param> -@ Acquisition - <1>" ("State")) -> (w4381:string)
        n1667 = call-poly <userlib>:"Build Message with Arguments++.vi"("States With Replace Token"=w4381, "<param>"=w4384, "<1>"=w4386) -> ("States"=w4385:string)  [unwired: 12 in]
        n1668 = in-place {
          in-place-border: w4379 -> [w4389]
          n1669 = in-place-cluster #41(w4380) -> ()  [unwired: 1 out]
          n1670 = in-place-cluster #41("Sample Settings.校准.校准模式"=w4389) -> (w4378:T20)
        }
        n1671 = call <vilib>:"Add State(s) to Queue__JKI_lib_State_Machine.vi"("State(s) in Front (\"\")"=w4385, "State(s) in (\"\")"=w4387) -> ("States Out"=w4388:string)  [unwired: 13 in]
      }
      frame "API: Dark Curnt Change" {
        n1672 = call "Convert API String Arguments to Data.vim"("Reference Type"=dbl[] [] ("温度校准值（每度）"), "API String"=w4396) -> ("Data"=w4395:dbl[])  [unwired: 6 in, 1 out]
        n1673 = Concatenate Strings(w4391, " >> <param> -@ Acquisition - <1>" ("State")) -> (w4390:string)
        n1674 = call-poly <userlib>:"Build Message with Arguments++.vi"("States With Replace Token"=w4390, "<param>"=w4396, "<1>"=w4398) -> ("States"=w4399:string)  [unwired: 12 in]
        n1675 = call <vilib>:"Add State(s) to Queue__JKI_lib_State_Machine.vi"("State(s) in Front (\"\")"=w4399, "State(s) in (\"\")"=w4400) -> ("States Out"=w4401:string)  [unwired: 13 in]
        n1676 = in-place {
          in-place-border: w4395 -> [w4403]
          n1677 = in-place-cluster #42(w4394) -> ()  [unwired: 1 out]
          n1678 = in-place-cluster #42("Sample Settings.校准.暗电流校准值初值"=w4403) -> (w4393:T20)
        }
      }
      frame "API: Dark Curnt Set to 0" {
        n1679 = Unbundle By Name(w4405) -> ("Sample Settings.设备信息.环数"=w4407:u8)
        n1680 = Initialize Array(0.0 ("暗电流校准值"), w4407) -> (w4406:dbl[])
        n1681 = local write "暗电流校准值"(w4406) -> ()
        n1682 = call "Convert Data To API String Arguments.vim"("Data"=w4406) -> ("API String"=w4412:string)  [unwired: 7 in, 1 out]
        n1683 = call-poly <userlib>:"Build Message with Arguments++.vi"("States With Replace Token"="API: Dark Curnt Change >> <param> -@ Acquisition - <1>" ("State"), "<param>"=w4412, "<1>"=w4409) -> ("States"=w4410:string)  [unwired: 12 in]
        n1684 = call <vilib>:"Add State(s) to Queue__JKI_lib_State_Machine.vi"("State(s) in Front (\"\")"=w4410, "State(s) in (\"\")"=w4413) -> ("States Out"=w4414:string)  [unwired: 13 in]
        n1685 = in-place {
          in-place-border: w4406 -> [w4416]
          n1686 = in-place-cluster #43(w4405) -> ()  [unwired: 1 out]
          n1687 = in-place-cluster #43("Sample Settings.校准.暗电流校准值初值"=w4416) -> (w4404:T20)
        }
      }
      frame "API: Wait" {
        n1688 = call "Convert API String Arguments to Data.vim"("Reference Type"=T14 {"每x周期/点等待"=0, "等待方式"=FALSE, "等待时间(s)"=0.0, "等待时"=enum."无电无光"} ("簇"), "API String"=w4428) -> ("Data"=w4423:T14)  [unwired: 6 in, 1 out]
        n1689 = Unbundle(w4423) -> ("每x周期/点等待"=w4421:i32, "等待方式"=w4420:bool, "等待时间(s)"=w4419:dbl, "等待时"=w4422:enum16{"无电无光", "有电无光", "无电有光", "有电有光"})
        n1690 = local write "等待时"(w4422) -> ()
        n1691 = local write "等待方式"(w4420) -> ()
        n1692 = local write "等待时间(s)"(w4419) -> ()
        n1693 = local write "每x周期/点等待"(w4421) -> ()
        n1694 = Concatenate Strings(w4426, " >> <param> -@ Acquisition - <1>" ("State")) -> (w4425:string)
        n1695 = call-poly <userlib>:"Build Message with Arguments++.vi"("States With Replace Token"=w4425, "<param>"=w4428, "<1>"=w4430) -> ("States"=w4429:string)  [unwired: 12 in]
        n1696 = in-place {
          in-place-border: w4422 -> [w4436]
          in-place-border: w4421 -> [w4433]
          in-place-border: w4420 -> [w4435]
          in-place-border: w4419 -> [w4434]
          n1697 = in-place-cluster #44(w4418) -> ()  [unwired: 4 out]
          n1698 = in-place-cluster #44("Sample Settings.等待.每x周期/点等待"=w4433, "Sample Settings.等待.等待方式"=w4435, "Sample Settings.等待.等待时间(s)"=w4434, "Sample Settings.等待.等待时"=w4436) -> (w4417:T20)
        }
        n1699 = call <vilib>:"Add State(s) to Queue__JKI_lib_State_Machine.vi"("State(s) in Front (\"\")"=w4429, "State(s) in (\"\")"=w4431) -> ("States Out"=w4432:string)  [unwired: 13 in]
      }
    }
  }
  n1700 = while {
    shift-right: [w4447] -> _
    shift-left: enum16{"Idle", "Initialize", "Exit"}."Initialize" -> [w4448]
    tunnel: "CSM Name" -> [w4445]
    shift-right: [w4443] -> _
    shift-left: w14 -> [w4444]
    shift-right: [w4441] -> _
    shift-left: -1 -> [w4442]
    shift-right: [w4440] -> _
    shift-left: _ -> [w4439]
    shift-right: [w4438] -> _
    shift-left: _ -> [w4437]
    stop <- w4446 stop-if-true
    n1701 = case shown="\"Idle\", 默认" w4448 {
      tunnel: [enum16{"Idle", "Initialize", "Exit"}."Idle" w4466 enum16{"Idle", "Initialize", "Exit"}."Exit"] -> w4447
      tunnel: [_ _ TRUE] -> w4446
      tunnel: w4445 -> [w4452 w4465 _]
      tunnel: w4444 -> [w4455 w4463 w4638]
      tunnel: [w4455 w4464 w4638] -> w4443
      tunnel: w4442 -> [_ w4461 _]
      tunnel: [-1 w4462 _] -> w4441
      tunnel: [w4451 w4459 _] -> w4440
      tunnel: w4439 -> [_ w4460 w4637]
      tunnel: [w4449 w4457 w4635] -> w4438
      tunnel: w4437 -> [_ w4458 w4635]
      frame "Initialize" {
        w4450 = FALSE  # your data
        n1702 = call <userlib>:"CSM - Module Exit Event.vi"("Name (\"\" to Use UUID) In"=w4452) -> ("CSM Exit Event"=w4453:refnum<user-event>)  [unwired: 8 in, 2 out]
        n1703 = register-events(w4453) -> (reference out=w4451:refnum<event-registration>)  [unwired: 2 in, 1 out]
        n1704 = Bundle("your data"=w4450) -> (w4449:cluster{"your data":bool})  [unwired: 1 in]
      }
      frame "Idle", Default {
        n1705 = event shown="[7] \"基准周期设定\": 值改变" {
          selector: w4460 -> [_ _ _ _ _ _ _ _ _ _ _ _ _ _ _ _ _ _ _ _ _ _ _ _]
          dyn-events: [_ _ _ _ _ _ _ _ _ _ _ _ _ _ _ _ _ _ _ _ _ _ _ _] -> w4459
          timeout: w4461 -> [_ _ _ _ _ _ _ _ _ _ _ _ _ _ _ _ _ _ _ _ _ _ _ _]
          tunnel: [_ w4473 enum16{"Idle", "Initialize", "Exit"}."Exit" _ _ _ _ _ _ _ _ _ _ _ _ _ _ _ _ _ _ _ _ _] -> w4466
          tunnel: w4465 -> [w4468 w4478 _ _ _ _ _ _ _ _ _ _ _ _ _ _ _ _ _ w4600 _ _ _ _]
          tunnel: w4463 -> [w4471 _ w4488 w4494 w4503 w4511 w4517 w4521 w4530 w4538 w4543 w4550 w4561 w4570 w4574 w4580 w4585 w4592 w4596 w4602 w4613 w4623 w4629 w4633]
          tunnel: [w4469 w4477 w4488 w4495 w4502 w4512 w4518 w4522 w4531 w4539 w4544 w4551 w4562 w4571 w4575 w4581 w4586 w4593 w4597 w4603 w4614 w4624 w4628 w4632] -> w4464
          tunnel: [-1 _ _ _ _ _ _ _ _ _ _ _ _ _ _ _ _ _ _ _ _ _ _ _] -> w4462
          tunnel: w4458 -> [w4467 w4476 w4486 w4496 w4504 w4515 w4519 w4523 w4532 w4540 w4547 w4554 w4565 w4572 w4576 w4583 w4587 w4594 w4598 w4604 w4615 w4626 w4630 w4634]
          tunnel: [w4467 w4476 w4486 w4496 w4504 w4515 w4519 w4523 w4532 w4540 w4547 w4554 w4565 w4572 w4576 w4583 w4587 w4594 w4598 w4604 w4615 w4626 w4630 w4634] -> w4457
          event Timeout {
            n1706 = event-data() -> ()  [unwired: 1 in, 3 out]
            n1707 = call-poly <userlib>:"CSM - Filter JKISM String Queue.vi"("States In"=w4471) -> ("States Out"=w4470:string)  [unwired: 14 in]
            n1708 = call <userlib>:"CSM - Forward UI Operations to CSM.vi"("Name (\"\" to Use UUID)"=w4468, "State(s) In (\"\")"=w4470) -> ("States Out"=w4469:string)  [unwired: 8 in, 1 out]
          }
          event Panel Close? {
            n1709 = event-data() -> ()  [unwired: 1 in, 1 out]
            n1710 = Two Button Dialog(message="确定关闭程序？" ("消息")) -> (T button?=w4474:bool)  [unwired: 2 in]
            n1711 = case shown="False" w4474 {
              tunnel: w4478 -> [w4481 w4484]
              tunnel: [w4481 w4483] -> w4477
              tunnel: [enum16{"Idle", "Initialize", "Exit"}."Idle" enum16{"Idle", "Initialize", "Exit"}."Exit"] -> w4473
              frame False {
              }
              frame True {
                n1712 = call <userlib>:"CSM - Forward UI Operations to CSM.vi"("Name (\"\" to Use UUID)"=w4484, "State(s) In (\"\")"="Macro: Exit" ("State")) -> ("States Out"=w4483:string)  [unwired: 8 in, 1 out]
              }
            }
            n1713 = event-data("Discard?"=TRUE) -> ()  [unwired: 1 in, 1 out]
          }
          event User Event {
            n1714 = event-data() -> ()  [unwired: 1 in, 1 out]
          }
          event "停止": Value Change {
            n1715 = event-data() -> ()  [unwired: 1 in, 1 out]
            n1716 = Two Button Dialog(message="确定停止程序？" ("消息")) -> (T button?=w4491:bool)  [unwired: 2 in]
            n1717 = Select(t="Macro: Exit" ("State(s) in Front (\"\")"), s=w4491, f="") -> (s? t:f=w4489:string)
            n1718 = call <vilib>:"Add State(s) to Queue__JKI_lib_State_Machine.vi"("State(s) in Front (\"\")"=w4489, "State(s) in (\"\")"=w4494) -> ("States Out"=w4495:string)  [unwired: 13 in]
          }
          event "开始": Value Change {
            n1719 = event-data() -> ()  [unwired: 1 in, 1 out]
            n1720 = flat-sequence {
              tunnel: [w4505] -> w4497
              frame #0 {
                n1721 = Two Button Dialog(message="是否追加数据？" ("消息"), 1:"否" ("F按钮名称（“取消”）"), 2:"是" ("T按钮名称（“确定”）")) -> (T button?=w4505:bool)
              }
            }
            n1722 = call "Convert Data To API String Arguments.vim"("Data"=w4497) -> ("API String"=w4500:string)  [unwired: 7 in, 1 out]
            n1723 = call <vilib>:"Build State String with Arguments__JKI_lib_State_Machine.vi"("Arguments (\"\")"=w4500, "State"="Macro: Start" ("State(s) in Front (\"\")")) -> ("State with Arguments"=w4498:string)  [unwired: 4 in]
            n1724 = local write "Error Occurred"(errorcluster {"status"=FALSE, "code"=0, "source"=""} ("错误常量")) -> ()
            n1725 = call <vilib>:"Add State(s) to Queue__JKI_lib_State_Machine.vi"("State(s) in Front (\"\")"=w4498, "State(s) in (\"\")"=w4503) -> ("States Out"=w4502:string)  [unwired: 13 in]
          }
          event "重新开始(不改变文件)": Value Change {
            n1726 = event-data() -> ()  [unwired: 1 in, 1 out]
            n1727 = call "Convert Data To API String Arguments.vim"("Data"=TRUE) -> ("API String"=w4514:string)  [unwired: 7 in, 1 out]
            n1728 = call <vilib>:"Build State String with Arguments__JKI_lib_State_Machine.vi"("Arguments (\"\")"=w4514, "State"="Macro: Start" ("State(s) in Front (\"\")")) -> ("State with Arguments"=w4510:string)  [unwired: 4 in]
            n1729 = call <vilib>:"Add State(s) to Queue__JKI_lib_State_Machine.vi"("State(s) in Front (\"\")"=w4510, "State(s) in (\"\")"=w4511) -> ("States Out"=w4512:string)  [unwired: 13 in]
          }
          event "暂停按钮": Value Change {
            n1730 = event-data() -> ()  [unwired: 1 in, 1 out]
            n1731 = call <vilib>:"Add State(s) to Queue__JKI_lib_State_Machine.vi"("State(s) in Front (\"\")"="Macro: Pause" ("State(s) in Front (\"\")"), "State(s) in (\"\")"=w4517) -> ("States Out"=w4518:string)  [unwired: 13 in]
          }
          event "基准周期设定": Value Change {
            n1732 = event-data() -> ()  [unwired: 1 in, 1 out]
            n1733 = call <vilib>:"Add State(s) to Queue__JKI_lib_State_Machine.vi"("State(s) in Front (\"\")"="Plot: Set Base Cycle to Current", "State(s) in (\"\")"=w4521) -> ("States Out"=w4522:string)  [unwired: 13 in]
          }
          event "测头拿取": Value Change {
            n1734 = event-data() -> ()  [unwired: 1 in, 1 out]
            n1735 = case shown="True" "计时方式" {
              frame False {
              }
              frame True {
                n1736 = local write "开始/清零"(FALSE ("暂停/继续")) -> ()
              }
            }
            n1737 = Select(t="API: Probe Up True", s="测头拿取", f="API: Probe Up False") -> (s? t:f=w4526:string)
            n1738 = Wait (ms)(milliseconds to wait=u32 100 ("等待时间（毫秒）")) -> ()  [unwired: 1 out]
            n1739 = call <vilib>:"Add State(s) to Queue__JKI_lib_State_Machine.vi"("State(s) in Front (\"\")"=w4526, "State(s) in (\"\")"=w4530) -> ("States Out"=w4531:string)  [unwired: 13 in]
          }
          event "测头供电": Value Change {
            n1740 = event-data() -> ()  [unwired: 1 in, 1 out]
            n1741 = call "Convert Data To API String Arguments.vim"("Data"="测头供电") -> ("API String"=w4536:string)  [unwired: 7 in, 1 out]
            n1742 = call <vilib>:"Build State String with Arguments__JKI_lib_State_Machine.vi"("Arguments (\"\")"=w4536, "State"="API: Probe Power") -> ("State with Arguments"=w4534:string)  [unwired: 4 in]
            n1743 = call <vilib>:"Add State(s) to Queue__JKI_lib_State_Machine.vi"("State(s) in Front (\"\")"=w4534, "State(s) in (\"\")"=w4538) -> ("States Out"=w4539:string)  [unwired: 13 in]
          }
          event "测头出光": Value Change {
            n1744 = event-data() -> ()  [unwired: 1 in, 1 out]
            n1745 = call "Convert Data To API String Arguments.vim"("Data"="测头出光") -> ("API String"=w4545:string)  [unwired: 7 in, 1 out]
            n1746 = call <vilib>:"Build State String with Arguments__JKI_lib_State_Machine.vi"("Arguments (\"\")"=w4545, "State"="API: Probe Light") -> ("State with Arguments"=w4542:string)  [unwired: 4 in]
            n1747 = call <vilib>:"Add State(s) to Queue__JKI_lib_State_Machine.vi"("State(s) in Front (\"\")"=w4542, "State(s) in (\"\")"=w4543) -> ("States Out"=w4544:string)  [unwired: 13 in]
          }
          event "是否保存": Value Change {
            n1748 = event-data() -> ()  [unwired: 1 in, 1 out]
            n1749 = call "Convert Data To API String Arguments.vim"("Data"="是否保存") -> ("API String"=w4552:string)  [unwired: 7 in, 1 out]
            n1750 = call <vilib>:"Build State String with Arguments__JKI_lib_State_Machine.vi"("Arguments (\"\")"=w4552, "State"="API: Data Save") -> ("State with Arguments"=w4549:string)  [unwired: 4 in]
            n1751 = call <vilib>:"Add State(s) to Queue__JKI_lib_State_Machine.vi"("State(s) in Front (\"\")"=w4549, "State(s) in (\"\")"=w4550) -> ("States Out"=w4551:string)  [unwired: 13 in]
          }
          event "等待方式", "等待时间(s)", "等待时", "每x周期/点等待": Value Change {
            n1752 = event-data() -> ()  [unwired: 1 in, 1 out]
            n1753 = Bundle("每x周期/点等待"="每x周期/点等待", "等待方式"="等待方式", "等待时间(s)"="等待时间(s)", "等待时"="等待时") -> (w4555:T22)  [unwired: 1 in]
            n1754 = call "Convert Data To API String Arguments.vim"("Data"=w4555) -> ("API String"=w4563:string)  [unwired: 7 in, 1 out]
            n1755 = call <vilib>:"Build State String with Arguments__JKI_lib_State_Machine.vi"("Arguments (\"\")"=w4563, "State"="API: Wait") -> ("State with Arguments"=w4560:string)  [unwired: 4 in]
            n1756 = call <vilib>:"Add State(s) to Queue__JKI_lib_State_Machine.vi"("State(s) in Front (\"\")"=w4560, "State(s) in (\"\")"=w4561) -> ("States Out"=w4562:string)  [unwired: 13 in]
          }
          event Value Change {
            n1757 = event-data() -> ()  [unwired: 1 in, 1 out]
            n1758 = call "Convert Data To API String Arguments.vim"("Data"="校准模式") -> ("API String"=w4568:string)  [unwired: 7 in, 1 out]
            n1759 = call <vilib>:"Build State String with Arguments__JKI_lib_State_Machine.vi"("Arguments (\"\")"=w4568, "State"="API: Dark Curnt Mode") -> ("State with Arguments"=w4567:string)  [unwired: 4 in]
            n1760 = call <vilib>:"Add State(s) to Queue__jki_lib_state_machine.vi"("State(s) in Front (\"\")"=w4567, "State(s) in (\"\")"=w4570) -> ("States Out"=w4571:string)  [unwired: 13 in]
          }
          event "暗电流赋0": Value Change {
            n1761 = event-data() -> ()  [unwired: 1 in, 1 out]
            n1762 = call <vilib>:"Add State(s) to Queue__JKI_lib_State_Machine.vi"("State(s) in Front (\"\")"="API: Dark Curnt Set to 0", "State(s) in (\"\")"=w4574) -> ("States Out"=w4575:string)  [unwired: 13 in]
          }
          event "暗电流校准值": Value Change {
            n1763 = event-data() -> ()  [unwired: 1 in, 1 out]
            n1764 = call "Convert Data To API String Arguments.vim"("Data"="暗电流校准值") -> ("API String"=w4577:string)  [unwired: 7 in, 1 out]
            n1765 = call <vilib>:"Build State String with Arguments__JKI_lib_State_Machine.vi"("Arguments (\"\")"=w4577, "State"="API: Dark Curnt Change") -> ("State with Arguments"=w4579:string)  [unwired: 4 in]
            n1766 = call <vilib>:"Add State(s) to Queue__JKI_lib_State_Machine.vi"("State(s) in Front (\"\")"=w4579, "State(s) in (\"\")"=w4580) -> ("States Out"=w4581:string)  [unwired: 13 in]
          }
          event "温度校准系数赋0": Value Change {
            n1767 = event-data() -> ()  [unwired: 1 in, 1 out]
            n1768 = call <vilib>:"Add State(s) to Queue__JKI_lib_State_Machine.vi"("State(s) in Front (\"\")"="Plot: Temp Calib Set to 0", "State(s) in (\"\")"=w4585) -> ("States Out"=w4586:string)  [unwired: 13 in]
          }
          event "温度校准值（每度）": Value Change {
            n1769 = event-data() -> ()  [unwired: 1 in, 1 out]
            n1770 = call "Convert Data To API String Arguments.vim"("Data"="温度校准值（每度）") -> ("API String"=w4591:string)  [unwired: 7 in, 1 out]
            n1771 = call <vilib>:"Build State String with Arguments__JKI_lib_State_Machine.vi"("Arguments (\"\")"=w4591, "State"="Plot: Temp Calib Change") -> ("State with Arguments"=w4588:string)  [unwired: 4 in]
            n1772 = call <vilib>:"Add State(s) to Queue__JKI_lib_State_Machine.vi"("State(s) in Front (\"\")"=w4588, "State(s) in (\"\")"=w4592) -> ("States Out"=w4593:string)  [unwired: 13 in]
          }
          event "图表重置": Value Change {
            n1773 = event-data() -> ()  [unwired: 1 in, 1 out]
            n1774 = call <vilib>:"Add State(s) to Queue__JKI_lib_State_Machine.vi"("State(s) in Front (\"\")"="Plot: Reset", "State(s) in (\"\")"=w4596) -> ("States Out"=w4597:string)  [unwired: 13 in]
          }
          event "分段颜色": Value Change {
            n1775 = event-data() -> ()  [unwired: 1 in, 1 out]
            n1776 = call "CSM Set Module Attribute.vim"("CSM Name"=w4600, "Attribute"="分段颜色", "Value"="分段颜色") -> ()  [unwired: 9 in, 4 out]
            n1777 = call <vilib>:"Add State(s) to Queue__JKI_lib_State_Machine.vi"("State(s) in (\"\")"=w4602) -> ("States Out"=w4603:string)  [unwired: 14 in]
          }
          event "单环上限", "单环下限", "单环图范围": Value Change {
            n1778 = event-data() -> ()  [unwired: 1 in, 1 out]
            n1779 = Bundle(cluster=T12 {"上限"=0.0, "下限"=0.0, "图范围"=enum."自动"} ("簇"), "上限"="单环上限", "下限"="单环下限", "图范围"="单环图范围") -> (w4608:T12)
            n1780 = call "Convert Data To API String Arguments.vim"("Data"=w4608) -> ("API String"=w4605:string)  [unwired: 7 in, 1 out]
            n1781 = call <vilib>:"Build State String with Arguments__JKI_lib_State_Machine.vi"("Arguments (\"\")"=w4605, "State"="Plot: sg_justify" ("消息")) -> ("State with Arguments"=w4606:string)  [unwired: 4 in]
            n1782 = call <vilib>:"Add State(s) to Queue__JKI_lib_State_Machine.vi"("State(s) in Front (\"\")"=w4606, "State(s) in (\"\")"=w4613) -> ("States Out"=w4614:string)  [unwired: 13 in]
          }
          event "差分上限", "差分下限", "差分图范围": Value Change {
            n1783 = event-data() -> ()  [unwired: 1 in, 1 out]
            n1784 = Bundle(cluster=T12 {"上限"=0.0, "下限"=0.0, "图范围"=enum."自动"} ("簇"), "上限"="差分上限", "下限"="差分下限", "图范围"="差分图范围") -> (w4621:T12)
            n1785 = call "Convert Data To API String Arguments.vim"("Data"=w4621) -> ("API String"=w4620:string)  [unwired: 7 in, 1 out]
            n1786 = call <vilib>:"Build State String with Arguments__JKI_lib_State_Machine.vi"("Arguments (\"\")"=w4620, "State"="Plot: diff_justify" ("消息")) -> ("State with Arguments"=w4622:string)  [unwired: 4 in]
            n1787 = call <vilib>:"Add State(s) to Queue__JKI_lib_State_Machine.vi"("State(s) in Front (\"\")"=w4622, "State(s) in (\"\")"=w4623) -> ("States Out"=w4624:string)  [unwired: 13 in]
          }
          event "添加": Value Change {
            n1788 = event-data() -> ()  [unwired: 1 in, 1 out]
            n1789 = call <vilib>:"Add State(s) to Queue__JKI_lib_State_Machine.vi"("State(s) in Front (\"\")"="Plot: Add Delta Curve" ("消息"), "State(s) in (\"\")"=w4629) -> ("States Out"=w4628:string)  [unwired: 13 in]
          }
          event "删除": Value Change {
            n1790 = event-data() -> ()  [unwired: 1 in, 1 out]
            n1791 = call <vilib>:"Add State(s) to Queue__JKI_lib_State_Machine.vi"("State(s) in Front (\"\")"="Plot: Delete Delta Curve" ("消息"), "State(s) in (\"\")"=w4633) -> ("States Out"=w4632:string)  [unwired: 13 in]
          }
        }
      }
      frame "Exit" {
        n1792 = Unregister For Events(event registration refnum=w4637) -> (error out=w4636:errorcluster)  [unwired: 1 in]
        n1793 = call <vilib>:"Clear Errors.vi"("error in (no error)"=w4636) -> ()  [unwired: 5 in, 2 out]
      }
    }
  }
  n1794 = flat-sequence {
    tunnel: w10 -> [_]
    tunnel: "CSM Name" -> [w4642]
    tunnel: "子程序？" -> [_]
    frame #0 {
      n1795 = Concatenate Strings("Acquisition - " ("Name(\"\" to use uuid)"), w4642) -> (w4644:string)
      n1796 = call "Acquisition.vi"("CSM Name"=w4644) -> ()  [unwired: 11 in]
      n1797 = Concatenate Strings("Logging - " ("Name(\"\" to use uuid)"), w4642) -> (w4641:string)
      n1798 = call "Logging.vi"("CSM Name"=w4641) -> ()  [unwired: 11 in]
    }
  }
  n1799 = Concatenate Strings("CSM Name", "_Time") -> (w2:string)
  n1800 = call <vilib>:"Add State(s) to Queue__JKI_lib_State_Machine.vi"("State(s) in (\"\")"="Macro: Initialize" ("Init State(\"Macro: Initialize\")")) -> ("States Out"=w4:string)  [unwired: 14 in]
  n1801 = while "Communicable State Machine(CSM) 2025" {
    shift-right: [w4660] -> _
    shift-left: _ -> [w4659]
    shift-right: [w4663] -> _
    shift-left: errorcluster {"status"=FALSE, "code"=0, "source"=""} ("error out") -> [w4657]
    shift-right: [w4662] -> _
    shift-left: w4 -> [w4664]
    tunnel: w2 -> [w4653]
    shift-right: [w4656] -> _
    shift-left: _ -> [w4647]
    shift-right: [w4655] -> _
    shift-left: _ -> [w4654]
    stop <- w4661 stop-if-true
    w4658 = -1  # Timeout
    # "#CSM Debug State History\n(delete if unneeded)"
    # "copy this to create labels for wires"
    # "System_Label"
    # "CSM Copyright ?2025 NEVSTOP https://github.com/NEVSTOP-LAB"
    n1802 = call <userlib>:"Parse State Queue++.vi"("State Queue"=w4664, "Name (\"\" to Use UUID)"=w4653, "Response Arguments"=w4647, "Previous Error"=w4657) -> ("Name Used"=w4648:string, "Remaining States"=w4665:string, "Current State"=w4652:string, "Arguments"=w4651:string, "Additional Information"=w4650:T15, "Source CSM"=w4649:string)  [unwired: 6 in]
    n1803 = call <userlib>:"CSM - Internal State Debug Log History.vi"("State"=w4652, "Arguments (\"\")"=w4651, ">> Response Source Message >>"=w4650, "Source (\"\")"=w4649) -> ("Debug Log"=→"State History - Time":string)  [unwired: 11 in]
    n1804 = case shown="\"UI: Initialize\"" w4652 {
      selector: w4652 -> [_ _ _ w4693 _ _ _ _ _ _ _ _ _ _ _ _ _ _ _ _ _ _ _ _ _ _ _ _ _ _ _]
      tunnel: w4665 -> [w4666 w4684 w4690 w4698 w4705 w4711 w4734 w4740 w4747 w4756 w4769 w4784 w4790 w4795 w4803 w4810 w4815 w4822 w4826 w4832 w4838 w4843 w4849 w4861 w4864 w4869 w4875 w4883 w4893 w4910 w4914]
      tunnel: w4651 -> [_ _ _ _ _ w4710 w4729 w4739 w4746 w4755 _ _ _ _ _ _ _ _ _ _ _ _ _ _ _ _ w4872 _ _ _ w4913]
      tunnel: w4659 -> [w4673 w4683 w4687 w4696 w4704 w4715 w4735 w4742 w4749 w4758 w4768 w4777 w4788 w4792 _ w4805 w4812 w4821 w4825 w4829 w4836 w4840 w4846 w4858 w4863 w4868 w4874 w4880 w4890 w4907 w4917]
      tunnel: [w4672 w4685 w4688 w4691 w4706 errorcluster {"status"=FALSE, "code"=0, "source"=""} ("error out") w4730 w4737 w4744 w4761 w4770 w4781 w4787 w4793 w4800 w4806 w4813 w4816 w4824 w4830 w4835 w4841 w4847 w4859 w4865 w4870 w4876 w4881 w4891 w4908 w4918] -> w4663
      tunnel: w4657 -> [w4671 w4685 w4688 w4699 w4706 w4712 w4736 w4738 w4745 _ w4770 w4781 w4787 w4793 w4800 w4807 w4813 _ w4827 w4830 w4835 w4841 w4847 w4859 w4865 w4870 w4876 w4881 w4891 w4908 w4918]
      tunnel: [w4674 w4684 w4689 w4697 w4705 w4707 w4733 w4743 w4750 w4757 w4769 w4783 w4789 w4794 w4802 w4809 w4814 w4822 w4826 w4831 w4837 w4842 w4848 w4860 w4864 w4869 w4875 w4882 w4892 w4909 w4915] -> w4662
      tunnel: [_ _ _ _ _ _ TRUE _ _ _ _ _ TRUE _ _ _ _ _ _ _ _ _ _ _ _ _ _ _ _ _ _] -> w4661
      tunnel: [w4670 w4683 w4687 w4696 w4704 w4715 w4735 w4742 w4749 w4759 w4768 w4782 w4788 w4792 w4801 w4805 w4812 w4821 w4825 w4829 w4836 w4840 w4846 w4858 w4863 w4868 w4874 w4880 w4890 w4907 w4917] -> w4660
      tunnel: w4658 -> [w4669 _ _ _ _ _ _ _ _ _ _ _ _ _ _ _ _ _ _ _ _ _ _ _ _ _ _ _ _ _ _]
      tunnel: w4649 -> [_ _ _ _ _ _ _ _ _ w4753 _ _ _ _ _ _ _ _ _ _ _ _ _ _ _ _ _ _ _ _ _]
      tunnel: w4650 -> [_ _ _ _ _ _ _ _ _ w4760 _ _ _ _ _ _ _ _ _ _ _ _ _ _ _ _ _ _ _ _ _]
      tunnel: [_ _ _ "" w4700 _ _ _ _ _ _ _ _ _ _ _ _ _ _ _ _ _ _ _ _ "API1 Response" w4871 _ _ _ _] -> w4656
      tunnel: [w4668 w4682 w4686 w4694 w4703 w4714 w4731 w4741 w4748 w4762 w4767 w4771 w4785 w4791 w4796 w4804 w4811 w4820 w4823 w4828 w4834 w4839 w4844 w4851 w4862 w4867 w4873 w4879 w4889 w4906 w4916] -> w4655
      tunnel: w4654 -> [w4668 w4682 w4686 w4694 w4703 w4714 w4731 w4741 w4748 w4762 w4767 w4771 w4785 w4791 w4796 w4804 w4811 _ w4823 w4828 w4834 w4839 w4844 w4851 w4862 w4867 w4873 w4879 w4889 w4906 w4916]
      tunnel: w4648 -> [_ _ _ w4692 _ _ w4728 _ _ _ _ _ _ _ _ _ _ w4819 _ _ _ _ _ _ _ _ _ _ _ _ _]
      frame "", "Event Structure", "Idle" {
        n1805 = call <userlib>:"Timeout Selector.vi"("Remaining States"=w4666, "Timeout Expected"=w4669) -> ("Timeout"=w4667:i32)  [unwired: 5 in]
        n1806 = event shown="[1] <New State Notifier Event>: 用户事件" {
          selector: w4668 -> [_ _]
          dyn-events: _ -> [_ _]
          timeout: w4667 -> [_ _]
          tunnel: w4666 -> [w4678 w4680]
          tunnel: [w4677 w4680] -> w4674
          tunnel: w4673 -> [w4675 w4681]
          tunnel: [w4676 w4679] -> w4672
          tunnel: w4671 -> [w4676 w4679]
          tunnel: [w4675 w4681] -> w4670
          event Timeout {
            n1807 = event-data() -> ()  [unwired: 1 in, 1 out]
            n1808 = call <vilib>:"Add State(s) to Queue__JKI_lib_State_Machine.vi"("State(s) in (\"\")"=w4678) -> ("States Out"=w4677:string)  [unwired: 14 in]
          }
          event User Event {
            # "#CSM \"New State Notifier Event\"\nThis user event is used to break out CSM from waiting in the event structure, to process the next state from external. DO NOT place any code here unless you really need to."
            n1809 = event-data() -> ()  [unwired: 1 in, 1 out]
          }
        }
      }
      frame "CSM Documentation" {
        # "#CSM README FIRST\n\nCommunicable State Machine(CSM) is a LabVIEW application framework that builds upon JKI State Machine(JKISM). It follows the pattern of JKISM and extends the keywords to describe message communication between modules, including concepts such as Sync-Message, Async-Message, Subscription/Unsubscription of status - essential elements for creating reusable code modules. For more information, please visit the CSM wiki: https://nevstop-lab.github.io/CSM-Wiki/\n\nFor instructions on JKI State Machine, visit: http://jki.net/state-machine/\nFor information about CSM, visit: https://github.com/NEVSTOP-LAB"
        # "#CSM \"Documentation\"\nCase for holding CSM Documenation"
      }
      frame "---------- Core ----------" {
        # "#CSM \"Category Seperator\"\nDo not put any code in this frame."
        n1810 = call <vilib>:"Add State(s) to Queue__JKI_lib_State_Machine.vi"("State(s) in (\"\")"=w4690) -> ("States Out"=w4689:string)  [unwired: 14 in]
      }
      frame Default {
        # "#CSM \"Default\"\nthis is used to capture unhandled states and typos"
        # "Handle mistyped state name (developer tool)"
        n1811 = call <userlib>:"CSM Unhandled State Error.vi"("error in (no error)"=w4699, "Undefined State"=w4693, "CSM Name"=w4692) -> ("error out"=w4691:errorcluster)  [unwired: 8 in]
        n1812 = call <vilib>:"Add State(s) to Queue__JKI_lib_State_Machine.vi"("State(s) in (\"\")"=w4698) -> ("States Out"=w4697:string)  [unwired: 14 in]
      }
      frame "VI Reference" {
        n1813 = Unbundle By Name(w4704) -> ("Core"=w4702:T16)
        n1814 = Unbundle By Name(w4702) -> ("Current VI Reference"=w4701:refnum<vi>)
        n1815 = call <userlib>:"CSM - Convert Data to HexStr.vi"("Variant"=w4701) -> ("HEX String (0-9,A-F)"=w4700:string)  [unwired: 8 in]
      }
      frame "Error Handler" {
        # "#CSM Disable this error dialog if you need"
        # "#CSM \"Error Handler\"\nYou can also output any states to clean-up after errors occur"
        # "Clear error"
        n1816 = case shown="错误" w4712 {
          selector: w4712 -> [_ w4722]
          tunnel: [w4721 w4724] -> w4708
          tunnel: w4711 -> [w4721 w4723]
          tunnel: w4710 -> [w4720 _]
          tunnel: [w4719 w4722] -> w4713
          frame No Error {
            n1817 = call <userlib>:"CSM - Convert Argument to Error.vi"("Argument"=w4720) -> ("Error"=w4719:errorcluster)  [unwired: 4 in]
            n1818 = flat-sequence {
              frame #0 {
                # "#CSM External Error Handler Case\nUsually, it's because This CSM register others' \"Error Occurred\" status with \"Error Handler\". If other CSM have any error, the error will be passed here for central handling."
              }
            }
          }
          frame Error {
            # "#CSM Internal Error Handler Case \nIf any error Occurred, \"Error Occurred\" \nstatus update will be broadcasted to system.\nParameter is Error Cluster."
            n1819 = call <userlib>:"CSM - Convert Error to Argument.vi"("Error"=w4722) -> ("Argument"=w4726:string)  [unwired: 4 in]
            n1820 = call <vilib>:"Build State String with Arguments__JKI_lib_State_Machine.vi"("Arguments (\"\")"=w4726, "State"="Error Occurred" ("Status with Arguments")) -> ("State with Arguments"=w4725:string)  [unwired: 4 in]
            n1821 = call <userlib>:"CSM - Broadcast Status Change.vi"("Status With Arguments"=w4725, "State Queue"=w4723) -> ("Remaining States"=w4724:string)  [unwired: 13 in]
          }
        }
        n1822 = disable-structure shown="Enabled" {
          disable-tunnel: w4713 -> [w4717 w4718]
          frame Enabled {
            n1823 = call <vilib>:"General Error Handler.vi"("error in (no error)"=w4717) -> ()  [unwired: 10 in, 5 out]
          }
          frame Disabled {
            n1824 = call <vilib>:"Clear Errors.vi"("error in (no error)"=w4718) -> ()  [unwired: 5 in, 2 out]
          }
        }
        n1825 = call <vilib>:"Add State(s) to Queue__JKI_lib_State_Machine.vi"("State(s) in Front (\"\")"="// Post Error States", "State(s) in (\"\")"=w4708) -> ("States Out"=w4707:string)  [unwired: 13 in]
      }
      frame "Critical Error" {
        # "#CSM Stop in Critical Error\nWhen Critical Error occurs, Stop the loop immediately. Do NOT change this unless you fully understand the impact."
        # "#CSM \"Critical Error\"\nWhen any un-recoverable error occurs, CSM goes into this case."
        n1826 = call <userlib>:"CSM Critical Error.vi"("error in (no error)"=w4736, "Arugments (As Reason)"=w4729, "CSM Name"=w4728) -> ("error out"=w4730:errorcluster)  [unwired: 8 in]
        n1827 = call <vilib>:"Add State(s) to Queue__JKI_lib_State_Machine.vi"("State(s) in (\"\")"=w4734) -> ("States Out"=w4733:string)  [unwired: 14 in]
      }
      frame "Target Error" {
        # "#CSM \"Target Error\"\nWhen This CSM try to communicate with an un-existed CSM, This CSM goes into this case."
        n1828 = call <userlib>:"CSM Target Error.vi"("error in (no error)"=w4738, "Arguments (As CSM Name)"=w4739) -> ("error out"=w4737:errorcluster)  [unwired: 9 in]
        n1829 = call <vilib>:"Add State(s) to Queue__JKI_lib_State_Machine.vi"("State(s) in (\"\")"=w4740) -> ("States Out"=w4743:string)  [unwired: 14 in]
      }
      frame "Target Timeout Error" {
        # "#CSM \"Target Timeout Error\"\nWhen This CSM could not get the sync-call response in time, This CSM goes into this case."
        n1830 = call <userlib>:"CSM Target Timeout Error.vi"("error in (no error)"=w4745, "Arguments (As CSM Name)"=w4746) -> ("error out"=w4744:errorcluster)  [unwired: 9 in]
        n1831 = call <vilib>:"Add State(s) to Queue__JKI_lib_State_Machine.vi"("State(s) in (\"\")"=w4747) -> ("States Out"=w4750:string)  [unwired: 14 in]
      }
      frame "Async Response", "Response" {
        n1832 = Unbundle(w4760) -> ("‘State"=w4754:string, "’Arguments"=w4752:string, "’Error"=w4751:errorcluster)
        n1833 = case shown="默认" w4754 {
          tunnel: [w4766] -> w4761
          tunnel: w4751 -> [w4766]
          tunnel: [w4765] -> w4759
          tunnel: w4758 -> [w4765]
          tunnel: [w4763] -> w4757
          tunnel: w4756 -> [w4764]
          tunnel: w4755 -> [_]
          tunnel: w4753 -> [_]
          tunnel: w4752 -> [_]
          frame 默认 {
            # "#CSM Response Comments\nAfter Message is executed, CSM goes to this state for receive the response.\n    For Async Message(->), \"Async Response\" is used. This CSM will goes to \"Async Message Posted\" immediately and receive the \"Async Response\" after the callee finishes the message.\n    For Sync Message(@),  This CSM will wait until the message is done and immediately goes to \"Response\""
            # "#CSM \"Async Response\"\nHandle Async-call Response (\"Async Response\" for ->)"
            # "#CSM \"Response\"\nHandle Sync-call Response (\"Response\" for -@)"
            n1834 = call <vilib>:"Add State(s) to Queue__JKI_lib_State_Machine.vi"("State(s) in (\"\")"=w4764) -> ("States Out"=w4763:string)  [unwired: 14 in]
          }
        }
      }
      frame "Async Message Posted" {
        # "#CSM \"Async Message Posted\"\nAfter Async Message is posted (-> or ->| ), CSM goes to this state for post-action.\nYou can use Argument - State to tell which Async Message is called."
      }
      frame "Initialize Core Data" {
        # "#CSM \"Initialize Core Data\"\nThis is used to determine panel behavior on exit"
        # "originally closed?"
        # "exe?"
        # "If panel starts closed or is an EXE, then close it when we exit"
        n1835 = property class="VI"() -> ("FP.State"=w4774:T9)  [unwired: 2 in, 2 out]
        n1836 = property class="App"() -> ("App.Kind"=w4780:T10)  [unwired: 2 in, 2 out]
        n1837 = control-ref of="Current VI Reference"() -> (w4775:refnum<vi>)
        n1838 = Equal?(x=w4774, y=T9."Closed" ("Front Panel Window:State")) -> (x = y?=w4772:bool)
        n1839 = Equal?(x=w4780, y=T10."Run Time System" ("Application:Kind")) -> (x = y?=w4778:bool)
        n1840 = Or(x=w4772, y=w4778) -> (x .or. y?=w4776:bool)
        n1841 = Bundle By Name(cluster=w4777, "Core.Current VI Reference"=w4775, "Core.Close Panel on Exit?"=w4776) -> (w4782:T23)
        n1842 = call <vilib>:"Add State(s) to Queue__JKI_lib_State_Machine.vi"("State(s) in (\"\")"=w4784) -> ("States Out"=w4783:string)  [unwired: 14 in]
      }
      frame "Exit" {
        # "#CSM \"Exit\"\nCase for exiting the loop. No errors that occur here will be handled."
        n1843 = call <vilib>:"Add State(s) to Queue__JKI_lib_State_Machine.vi"("State(s) in (\"\")"=w4790) -> ("States Out"=w4789:string)  [unwired: 14 in]
      }
      frame "---------- Data ----------" {
        # "#CSM \"Category Seperator\"\nDo not put any code in this frame."
        n1844 = call <vilib>:"Add State(s) to Queue__JKI_lib_State_Machine.vi"("State(s) in (\"\")"=w4795) -> ("States Out"=w4794:string)  [unwired: 14 in]
      }
      frame "Data: Initialize" {
        w4797 = T16 {"Current VI Reference"=refnum, "Close Panel on Exit?"=FALSE}  # Core
        w4799 = TRUE  # Your Boolean data
        w4798 = ""  # Your string data
        # "#CSM do not delete - used by framework"
        # "#CSM Expand Bundle to add new data elements to shift register data."
        # "#CSM Add new data here."
        # "Initialize the shift-register data, here.\n(data names are defined by what you wire into the bundle function)"
        n1845 = Bundle("Core"=w4797, "Your Boolean data"=w4799, "Your string data"=w4798) -> (w4801:T23)  [unwired: 1 in]
        n1846 = call <vilib>:"Add State(s) to Queue__JKI_lib_State_Machine.vi"("State(s) in (\"\")"=w4803) -> ("States Out"=w4802:string)  [unwired: 14 in]
      }
      frame "Data: Cleanup" {
        # "Cleanup any data and references, here.\n(this is called automatically, by the Macro: Exit)"
        n1847 = Unbundle By Name(w4805) -> ("Core.Current VI Reference"=w4808:refnum<vi>)
        n1848 = Close Reference(reference=w4808, error in (no error)=w4807) -> (error out=w4806:errorcluster)
        n1849 = call <vilib>:"Add State(s) to Queue__JKI_lib_State_Machine.vi"("State(s) in (\"\")"=w4810) -> ("States Out"=w4809:string)  [unwired: 14 in]
      }
      frame "---------- Events ----------" {
        # "#CSM \"Category Seperator\"\nDo not put any code in this frame."
        n1850 = call <vilib>:"Add State(s) to Queue__JKI_lib_State_Machine.vi"("State(s) in (\"\")"=w4815) -> ("States Out"=w4814:string)  [unwired: 14 in]
      }
      frame "Events: Register" {
        # "#CSM \"Events: Register\"\nRegister user event. New Message Event is registered to break CSM waiting in event structure by default."
        # "#CSM Register New Message Event\nRegister message event to break Waiting in Event structure."
        n1851 = call <userlib>:"CSM - Get New State Notifier Event.vi"("Name (\"\" to Use UUID)"=w4819) -> ("error out"=w4817:errorcluster, "New State Notifier Event"=w4818:refnum<user-event>)  [unwired: 9 in]
        n1852 = register-events(error in=w4817, w4818) -> (reference out=w4820:refnum<event-registration>, error out=w4816:errorcluster)  [unwired: 1 in]
      }
      frame "Events: Unregister" {
        # "#CSM \"Events: Unregister\"\nUnregister user event."
        n1853 = Unregister For Events(event registration refnum=w4823, error in=w4827) -> (error out=w4824:errorcluster)
      }
      frame "---------- UI ----------" {
        # "#CSM \"Category Seperator\"\nDo not put any code in this frame."
        n1854 = call <vilib>:"Add State(s) to Queue__JKI_lib_State_Machine.vi"("State(s) in (\"\")"=w4832) -> ("States Out"=w4831:string)  [unwired: 14 in]
      }
      frame "UI: Initialize" {
        # "#CSM \"UI: Initialize\"\nInitialize the User Interface, here.\n(this is called automatically, by the Macro: Init)"
        n1855 = local write "开始/清零"(FALSE ("开始/清零")) -> ()
        n1856 = call <vilib>:"Add State(s) to Queue__JKI_lib_State_Machine.vi"("State(s) in (\"\")"=w4838) -> ("States Out"=w4837:string)  [unwired: 14 in]
      }
      frame "---------- Macro ----------" {
        # "#CSM \"Category Seperator\"\nDo not put any code in this frame."
        n1857 = call <vilib>:"Add State(s) to Queue__JKI_lib_State_Machine.vi"("State(s) in (\"\")"=w4843) -> ("States Out"=w4842:string)  [unwired: 14 in]
      }
      frame "Macro: Initialize" {
        # "#CSM \"Macro: Initialize\"\nInitialization Macro (This is called once, when the VI starts)"
        n1858 = call <vilib>:"Add State(s) to Queue__JKI_lib_State_Machine.vi"("State(s) in Front (\"\")"="Data: Initialize\nInitialize Core Data\nEvents: Register\nUI: Initialize\n\nTime: Sys Time", "State(s) in (\"\")"=w4849) -> ("States Out"=w4848:string)  [unwired: 13 in]
      }
      frame "Macro: Exit" {
        # "#CSM \"Macro: Exit\"\nExit Macro (This is called once, when the VI exits)"
        n1859 = Unbundle By Name(w4858) -> ("Core.Close Panel on Exit?"=w4857:bool)
        n1860 = Select(t="UI: Front Panel State >> Close", s=w4857, f="") -> (s? t:f=w4854:string)
        n1861 = call <vilib>:"Add State(s) to Queue__JKI_lib_State_Machine.vi"("State(s) in Front (\"\")"="//Exit Sub-Modules ", "State(s) in (\"\")"=w4854, "State(s) at Back (\"\")"="Data: Cleanup\nEvents: Unregister\nExit") -> ("States Out"=w4852:string)  [unwired: 12 in]
        n1862 = call <vilib>:"Add State(s) to Queue__JKI_lib_State_Machine.vi"("State(s) in Front (\"\")"=w4852, "State(s) in (\"\")"=w4861) -> ("States Out"=w4860:string)  [unwired: 13 in]
      }
      frame "---------- API ----------" {
        # "#CSM \"Category Seperator\"\nDo not put any code in this frame."
      }
      frame "API: API1" {
        # "#CSM API Example\nCopy/Rename this case for your own API"
        # "#CSM Response\nConnect this to return the response of your API"
        # "#CSM >> Source CSM >>\nIf you need to tell who triggered this state , use this string. If it's this case itself, this string is \"\"."
        # "#CSM >> Arguments >>\nDeal with the parameter if any"
      }
      frame "API: API2" {
        # "#CSM API Example\nCopy/Rename this case for your own API"
        # "unpack Hex String  to Variant\nif complex parameter is needed."
        n1863 = call <userlib>:"CSM - Convert HexStr to Data.vi"("HEX String"=w4872) -> ()  [unwired: 7 in, 2 out]
        n1864 = disable-structure shown="Disabled" {
          disable-tunnel: [w4877 "API2 Response"] -> w4871
          frame Disabled {
            # "pack variant to hexstr \nif complex response is needed."
            # "complex Response"
            n1865 = call <userlib>:"CSM - Convert Data to HexStr.vi"() -> ("HEX String (0-9,A-F)"=w4877:string)  [unwired: 9 in]
          }
          frame Enabled {
          }
        }
      }
      frame "---------- Time ----------" {
        # "#CSM \"Category Seperator\"\nDo not put any code in this frame."
        n1866 = call <vilib>:"Add State(s) to Queue__JKI_lib_State_Machine.vi"("State(s) in (\"\")"=w4883) -> ("States Out"=w4882:string)  [unwired: 14 in]
      }
      frame "Time: Sys Time" {
        # "#CSM \"Internal State\"\nThis category is used for holding internal states"
        n1867 = Get Date/Time In Seconds() -> (seconds since 1Jan1904=w4888:timestamp)
        n1868 = Format Date/Time String(time format string (%c)="%H: %M: %S" ("时间格式字符串(%c)"), seconds (now)=w4888) -> (date/time string=→"时间":string)  [unwired: 1 in]
        n1869 = Wait (ms)(milliseconds to wait=u32 50 ("等待时间（毫秒）")) -> ()  [unwired: 1 out]
        n1870 = call <vilib>:"Add State(s) to Queue__JKI_lib_State_Machine.vi"("State(s) in (\"\")"=w4893, "State(s) at Back (\"\")"="Time: Meas Time\nTime: Sys Time") -> ("States Out"=w4892:string)  [unwired: 13 in]
      }
      frame "Time: Meas Time" {
        # "start\n拿起\n放下"
        # "#CSM \"Internal State\"\nThis category is used for holding internal states"
        n1871 = Select(t=enum16{"开始计时", "暂停", "继续"}."继续" ("动作"), s="暂停/继续", f=enum16{"开始计时", "暂停", "继续"}."暂停") -> (s? t:f=w4900:enum16{"开始计时", "暂停", "继续"})
        n1872 = Select(t=w4900, s="开始/清零", f=enum16{"开始计时", "暂停", "继续"}."开始计时") -> (s? t:f=w4901:enum16{"开始计时", "暂停", "继续"})
        n1873 = Wait (ms)(milliseconds to wait=u32 50 ("等待时间（毫秒）")) -> ()  [unwired: 1 out]
        n1874 = call "FGV_new.vi"("动作"=w4901) -> ("计时时间"=w4905:dbl)  [unwired: 8 in, 2 out]
        n1875 = Format Date/Time String(time format string (%c)="%H: %M: %S" ("时间格式字符串(%c)"), seconds (now)=w4905, UTC format=TRUE ("UTC格式")) -> (date/time string=→"计时":string)
        n1876 = call <vilib>:"Add State(s) to Queue__JKI_lib_State_Machine.vi"("State(s) in (\"\")"=w4910) -> ("States Out"=w4909:string)  [unwired: 14 in]
      }
      frame "Time: Wait Count" {
        n1877 = call "Convert API String Arguments to Data.vim"("Reference Type"=0.0 ("下限"), "API String"=w4913) -> ("Data"=→"等待倒计时(s)":dbl)  [unwired: 6 in, 1 out]
        n1878 = call <vilib>:"Add State(s) to Queue__JKI_lib_State_Machine.vi"("State(s) in (\"\")"=w4914) -> ("States Out"=w4915:string)  [unwired: 14 in]
      }
    }
  }
  n1879 = call <userlib>:"CSM - Sync Configuration Variables to File.vi"("All Temp Variable to Default Ini(F)"=TRUE, "error in (no error)"=w8) -> ()  [unwired: 7 in, 1 out]
